vi "Edit Curve.vi"(8 "error in (no error)":errorcluster, 10 "Plot Index":i32, 11 "Data Viewer in":refnum<class "Data Viewer.lvclass">) -> (0 "error out":errorcluster, 1 "Cancel?":bool, 3 "Data Viewer out":refnum<class "Data Viewer.lvclass">)   [LabVIEW 2020, in "Data Viewer.lvlib" / "Data Viewer.lvclass"]
uses:
  Data Viewer.lvclass
  Data Viewer.lvclass/Data Viewer.ctl
panel:
  in  "Tab Control":enum32{"Page 2"}(tab)
  out "名称":string
  in  "Accept":bool
  in  "Data Array":cluster{"Time":timestamp, "Value":dbl}[](array[cluster]) {"Value" format="%.3f"; "Time" format="%<%Y/%m/%d %H:%M:%S%3u>T"}
  in  "Date":timestamp format="%<%Y/%m/%d %H:%M:%S%3u>T"
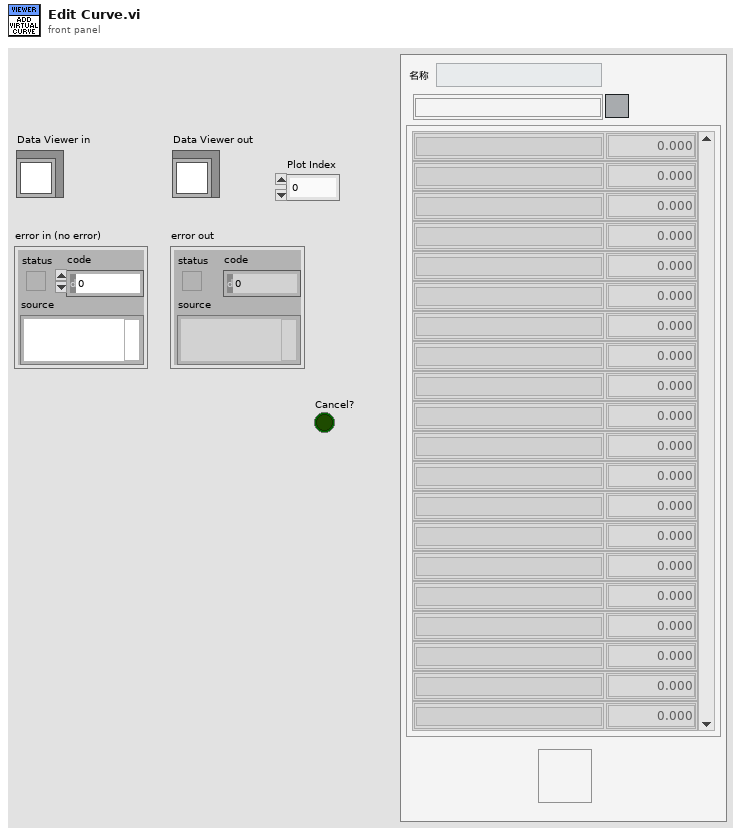
[diagram p1: front panel]
types:
  T1 = enum32{"Invalid", "Standard", "Closed", "Hidden", "Minimized", "Maximized"}
  T2 = typedef "Data Viewer.lvlib/Data Viewer.lvclass/Plot Property--cluster.ctl" = cluster{"Name":string, "Visible":bool, "Color":u32, "Scale Index":i32, "Show Peak Line":bool}
  T3 = typedef "Data Viewer.lvlib/Data Serie--cluster.ctl" = cluster{"Name":string, "Unit":string, "Sample Rate[Hz]":dbl, "Delta t[S]":dbl, "t0":timestamp, "Length":i32, "Time":timestamp[], "Value":dbl[]}
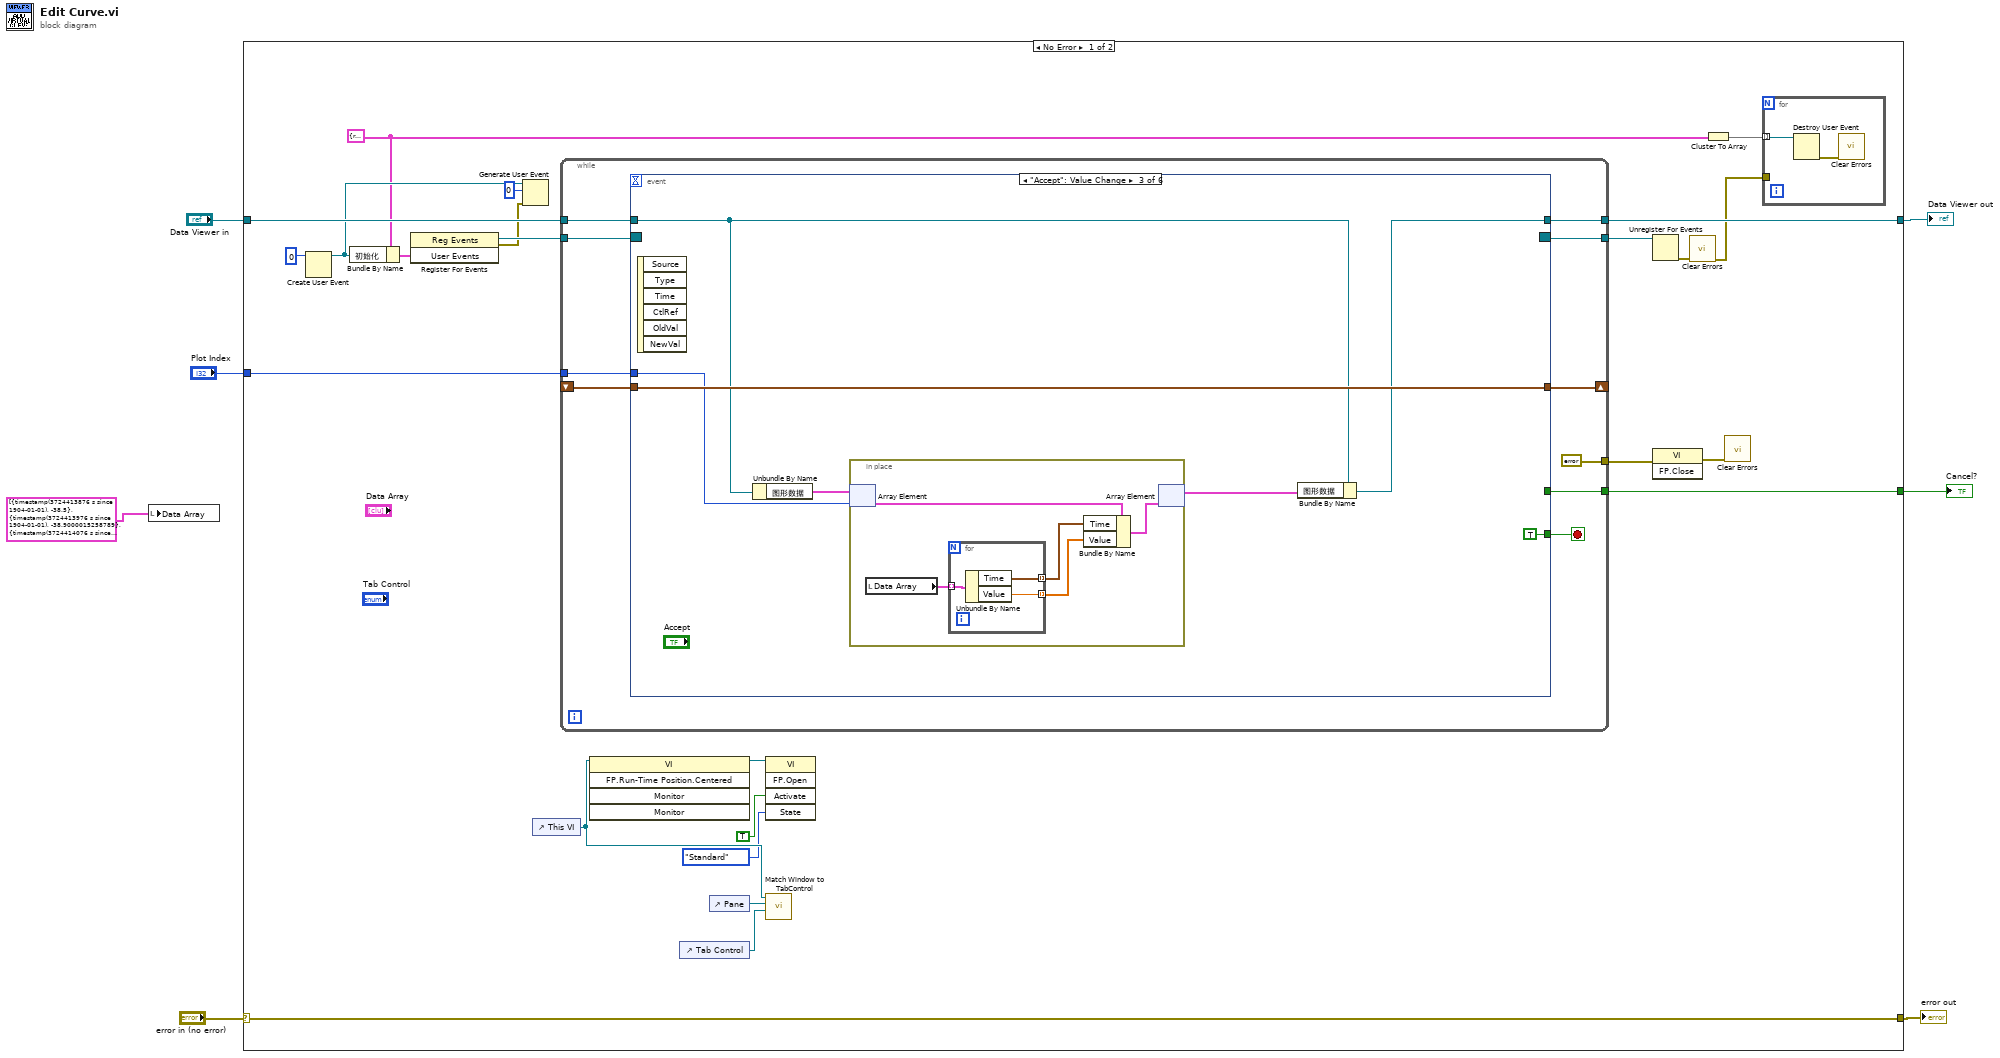
[diagram p0: block diagram]
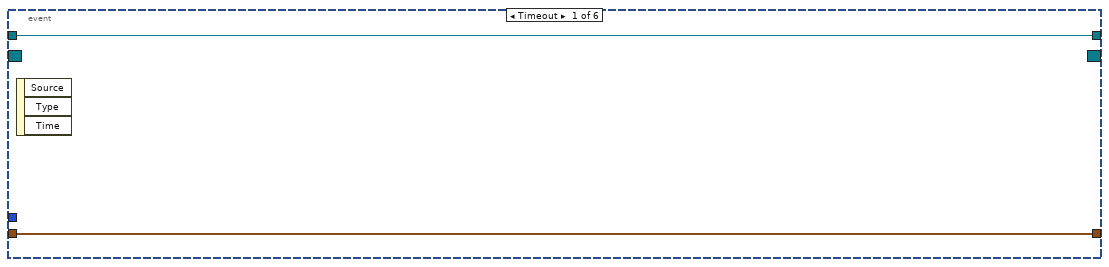
[diagram p2: hidden frame]
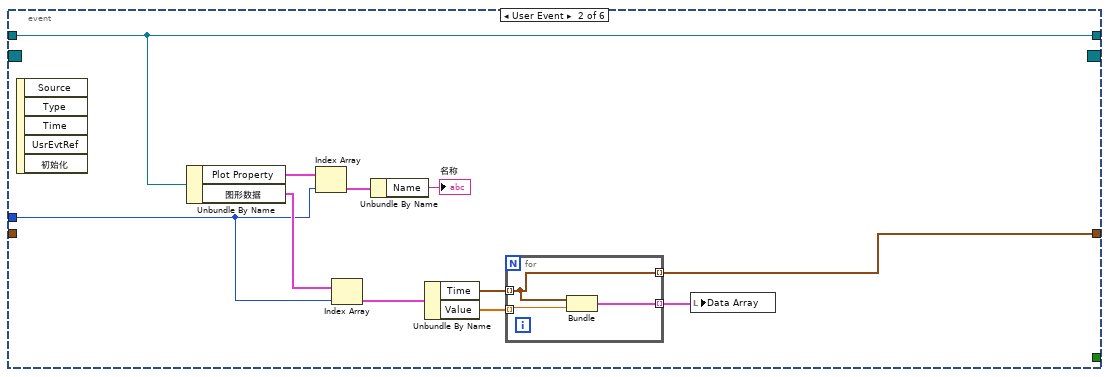
[diagram p3: hidden frame]
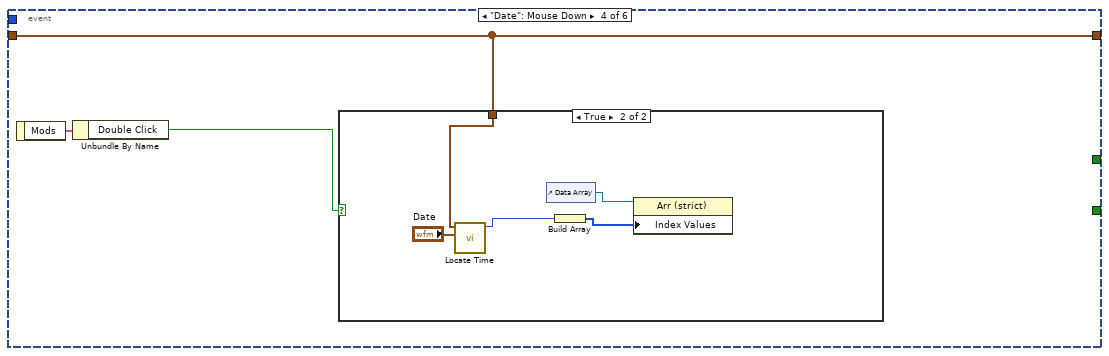
[diagram p4: hidden frame]
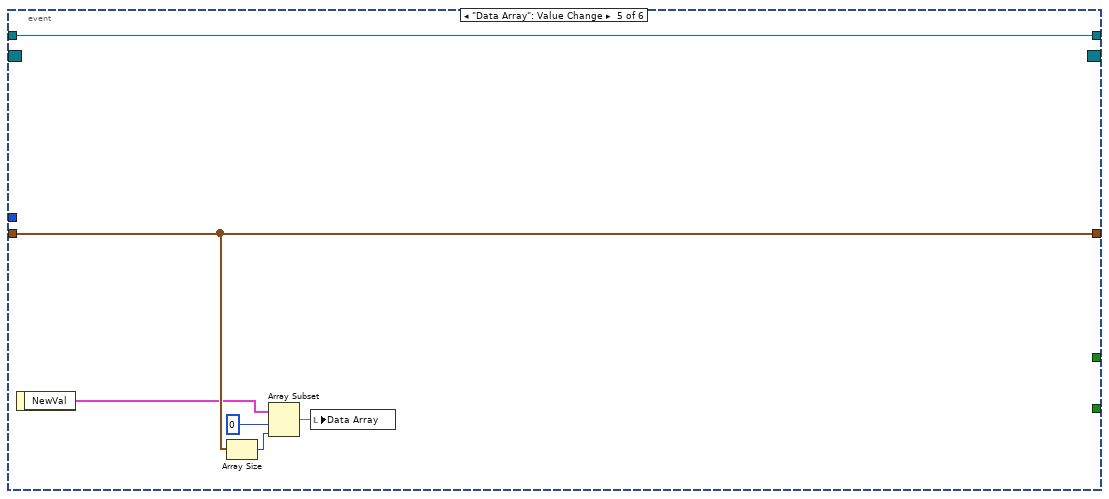
[diagram p6: hidden frame]
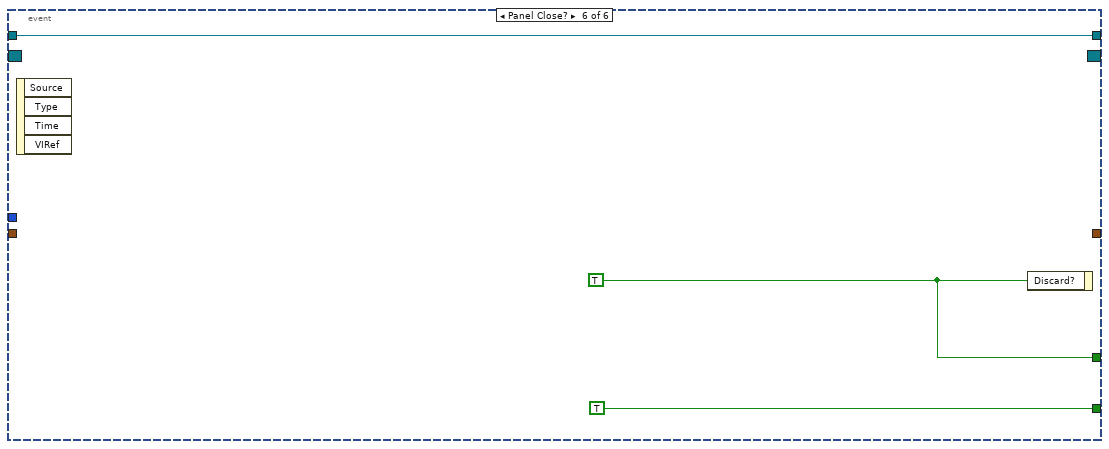
[diagram p7: hidden frame]
diagram:
  n1 = local write "Data Array"(cluster{"数值":timestamp, "数值 2":dbl}[] [{"数值"=timestamp(3724413876.000003 s since 1904-01-01), "数值 2"=-38.5}, {"数值"=timestamp(3724413976.000003 s since 1904-01-01), "数值 2"=-38.9000015258789}, {"数值"=timestamp(3724414076.000003 s since 1904-01-01), "数值 2"=-40.7000007629395}, {"数值"=timestamp(3724414176.000003 s since 1904-01-01), "数值 2"=-41.2000007629395}, {"数值"=timestamp(3724414276.000003 s since 1904-01-01), "数值 2"=-40.5999984741211}, {"数值"=timestamp(3724414376.000003 s since 1904-01-01), "数值 2"=-38.7000007629395}, {"数值"=timestamp(3724414476.000003 s since 1904-01-01), "数值 2"=-38.7000007629395}, {"数值"=timestamp(3724414576.000003 s since 1904-01-01), "数值 2"=-40.4000015258789}, {"数值"=timestamp(3724414676.000003 s since 1904-01-01), "数值 2"=-41.0999984741211}, {"数值"=timestamp(3724414776.000003 s since 1904-01-01), "数值 2"=-40.7999992370605}, {"数值"=timestamp(3724414876.000003 s since 1904-01-01), "数值 2"=-39.5999984741211}, {"数值"=timestamp(3724414976.000003 s since 1904-01-01), "数值 2"=59.5}, {"数值"=timestamp(3724415076.000003 s since 1904-01-01), "数值 2"=86.3000030517578}, {"数值"=timestamp(3724415176.000003 s since 1904-01-01), "数值 2"=85.1999969482422}, {"数值"=timestamp(3724415276.000003 s since 1904-01-01), "数值 2"=85.0999984741211}, {"数值"=timestamp(3724415376.000003 s since 1904-01-01), "数值 2"=85.0}, {"数值"=timestamp(3724415476.000003 s since 1904-01-01), "数值 2"=85.0}, {"数值"=timestamp(3724415576.000003 s since 1904-01-01), "数值 2"=85.0}, {"数值"=timestamp(3724415676.000003 s since 1904-01-01), "数值 2"=85.0}, {"数值"=timestamp(3724415776.000003 s since 1904-01-01), "数值 2"=85.0}, {"数值"=timestamp(3724415876.000003 s since 1904-01-01), "数值 2"=85.0}, {"数值"=timestamp(3724415976.000003 s since 1904-01-01), "数值 2"=85.0}, {"数值"=timestamp(3724416076.000003 s since 1904-01-01), "数值 2"=85.0}, {"数值"=timestamp(3724416176.000003 s since 1904-01-01), "数值 2"=85.0999984741211}, {"数值"=timestamp(3724416276.000003 s since 1904-01-01), "数值 2"=84.9000015258789}, {"数值"=timestamp(3724416376.000003 s since 1904-01-01), "数值 2"=84.9000015258789}, {"数值"=timestamp(3724416476.000003 s since 1904-01-01), "数值 2"=84.9000015258789}, {"数值"=timestamp(3724416576.000003 s since 1904-01-01), "数值 2"=85.0}, {"数值"=timestamp(3724416676.000003 s since 1904-01-01), "数值 2"=85.0}, {"数值"=timestamp(3724416776.000003 s since 1904-01-01), "数值 2"=-2.0}, {"数值"=timestamp(3724416876.000003 s since 1904-01-01), "数值 2"=-42.5}, {"数值"=timestamp(3724416976.000003 s since 1904-01-01), "数值 2"=-40.7999992370605}, {"数值"=timestamp(3724417076.000003 s since 1904-01-01), "数值 2"=-40.2999992370605}, {"数值"=timestamp(3724417176.000003 s since 1904-01-01), "数值 2"=-38.0999984741211}, {"数值"=timestamp(3724417276.000003 s since 1904-01-01), "数值 2"=-38.2000007629395}, {"数值"=timestamp(3724417376.000003 s since 1904-01-01), "数值 2"=-39.0999984741211}, {"数值"=timestamp(3724417476.000003 s since 1904-01-01), "数值 2"=-40.4000015258789}, {"数值"=timestamp(3724417576.000003 s since 1904-01-01), "数值 2"=-41.0}, {"数值"=timestamp(3724417676.000003 s since 1904-01-01), "数值 2"=-41.0}, {"数值"=timestamp(3724417776.000003 s since 1904-01-01), "数值 2"=-39.7000007629395}, {"数值"=timestamp(3724417876.000003 s since 1904-01-01), "数值 2"=-38.5999984741211}, {"数值"=timestamp(3724417976.000003 s since 1904-01-01), "数值 2"=-39.2999992370605}, {"数值"=timestamp(3724418076.000003 s since 1904-01-01), "数值 2"=-40.9000015258789}, {"数值"=timestamp(3724418176.000003 s since 1904-01-01), "数值 2"=-41.2000007629395}, {"数值"=timestamp(3724418276.000003 s since 1904-01-01), "数值 2"=-40.5999984741211}, {"数值"=timestamp(3724418376.000003 s since 1904-01-01), "数值 2"=-38.7999992370605}, {"数值"=timestamp(3724418476.000003 s since 1904-01-01), "数值 2"=-38.5999984741211}, {"数值"=timestamp(3724418576.000003 s since 1904-01-01), "数值 2"=-40.0999984741211}, {"数值"=timestamp(3724418676.000003 s since 1904-01-01), "数值 2"=-41.0999984741211}, {"数值"=timestamp(3724418776.000003 s since 1904-01-01), "数值 2"=-40.9000015258789}, {"数值"=timestamp(3724418876.000003 s since 1904-01-01), "数值 2"=-39.9000015258789}, {"数值"=timestamp(3724418976.000003 s since 1904-01-01), "数值 2"=-38.5999984741211}, {"数值"=timestamp(3724419076.000003 s since 1904-01-01), "数值 2"=-39.5999984741211}, {"数值"=timestamp(3724419176.000003 s since 1904-01-01), "数值 2"=-40.7000007629395}, {"数值"=timestamp(3724419276.000003 s since 1904-01-01), "数值 2"=-41.0999984741211}, {"数值"=timestamp(3724419376.000003 s since 1904-01-01), "数值 2"=-40.4000015258789}, {"数值"=timestamp(3724419476.000003 s since 1904-01-01), "数值 2"=-37.0}, {"数值"=timestamp(3724419576.000003 s since 1904-01-01), "数值 2"=86.4000015258789}, {"数值"=timestamp(3724419676.000003 s since 1904-01-01), "数值 2"=85.0}, {"数值"=timestamp(3724419776.000003 s since 1904-01-01), "数值 2"=85.0999984741211}, {"数值"=timestamp(3724419876.000003 s since 1904-01-01), "数值 2"=85.0}, {"数值"=timestamp(3724419976.000003 s since 1904-01-01), "数值 2"=84.9000015258789}, {"数值"=timestamp(3724420076.000003 s since 1904-01-01), "数值 2"=84.9000015258789}, {"数值"=timestamp(3724420176.000003 s since 1904-01-01), "数值 2"=85.0}, {"数值"=timestamp(3724420276.000003 s since 1904-01-01), "数值 2"=85.0}, {"数值"=timestamp(3724420376.000003 s since 1904-01-01), "数值 2"=85.0999984741211}, {"数值"=timestamp(3724420476.000003 s since 1904-01-01), "数值 2"=84.9000015258789}, {"数值"=timestamp(3724420576.000003 s since 1904-01-01), "数值 2"=84.9000015258789}, {"数值"=timestamp(3724420676.000003 s since 1904-01-01), "数值 2"=85.0}, {"数值"=timestamp(3724420776.000003 s since 1904-01-01), "数值 2"=85.0}, {"数值"=timestamp(3724420876.000003 s since 1904-01-01), "数值 2"=85.0}, {"数值"=timestamp(3724420976.000003 s since 1904-01-01), "数值 2"=84.9000015258789}, {"数值"=timestamp(3724421076.000003 s since 1904-01-01), "数值 2"=85.0999984741211}, {"数值"=timestamp(3724421176.000003 s since 1904-01-01), "数值 2"=85.0}, {"数值"=timestamp(3724421276.000003 s since 1904-01-01), "数值 2"=76.1999969482422}, {"数值"=timestamp(3724421376.000003 s since 1904-01-01), "数值 2"=-42.0999984741211}, {"数值"=timestamp(3724421476.000003 s since 1904-01-01), "数值 2"=-40.7999992370605}, {"数值"=timestamp(3724421576.000003 s since 1904-01-01), "数值 2"=-40.2999992370605}, {"数值"=timestamp(3724421676.000003 s since 1904-01-01), "数值 2"=-38.0}, {"数值"=timestamp(3724421776.000003 s since 1904-01-01), "数值 2"=-38.2999992370605}, {"数值"=timestamp(3724421876.000003 s since 1904-01-01), "数值 2"=-39.0999984741211}, {"数值"=timestamp(3724421976.000003 s since 1904-01-01), "数值 2"=-40.7000007629395}, {"数值"=timestamp(3724422076.000003 s since 1904-01-01), "数值 2"=-41.2000007629395}, {"数值"=timestamp(3724422176.000003 s since 1904-01-01), "数值 2"=-40.9000015258789}, {"数值"=timestamp(3724422276.000003 s since 1904-01-01), "数值 2"=-39.2999992370605}, {"数值"=timestamp(3724422376.000003 s since 1904-01-01), "数值 2"=-38.7000007629395}, {"数值"=timestamp(3724422476.000003 s since 1904-01-01), "数值 2"=-39.9000015258789}, {"数值"=timestamp(3724422576.000003 s since 1904-01-01), "数值 2"=-41.0}, {"数值"=timestamp(3724422676.000003 s since 1904-01-01), "数值 2"=-41.0}, {"数值"=timestamp(3724422776.000003 s since 1904-01-01), "数值 2"=-40.2000007629395}, {"数值"=timestamp(3724422876.000003 s since 1904-01-01), "数值 2"=-38.5999984741211}, {"数值"=timestamp(3724422976.000003 s since 1904-01-01), "数值 2"=-39.0}, {"数值"=timestamp(3724423076.000003 s since 1904-01-01), "数值 2"=-40.5}, {"数值"=timestamp(3724423176.000003 s since 1904-01-01), "数值 2"=-41.2000007629395}, {"数值"=timestamp(3724423276.000003 s since 1904-01-01), "数值 2"=-40.7999992370605}, {"数值"=timestamp(3724423376.000003 s since 1904-01-01), "数值 2"=-39.5999984741211}, {"数值"=timestamp(3724423476.000003 s since 1904-01-01), "数值 2"=-38.5999984741211}, {"数值"=timestamp(3724423576.000003 s since 1904-01-01), "数值 2"=-39.7999992370605}, {"数值"=timestamp(3724423676.000003 s since 1904-01-01), "数值 2"=-40.7999992370605}, {"数值"=timestamp(3724423776.000003 s since 1904-01-01), "数值 2"=-41.0}, {"数值"=timestamp(3724423876.000003 s since 1904-01-01), "数值 2"=-40.2000007629395}, {"数值"=timestamp(3724423976.000003 s since 1904-01-01), "数值 2"=-6.90000009536743}, {"数值"=timestamp(3724424076.000003 s since 1904-01-01), "数值 2"=86.0}, {"数值"=timestamp(3724424176.000003 s since 1904-01-01), "数值 2"=85.0999984741211}, {"数值"=timestamp(3724424276.000003 s since 1904-01-01), "数值 2"=85.0}, {"数值"=timestamp(3724424376.000003 s since 1904-01-01), "数值 2"=85.0}, {"数值"=timestamp(3724424476.000003 s since 1904-01-01), "数值 2"=85.0}, {"数值"=timestamp(3724424576.000003 s since 1904-01-01), "数值 2"=85.0}, {"数值"=timestamp(3724424676.000003 s since 1904-01-01), "数值 2"=85.0}, {"数值"=timestamp(3724424776.000003 s since 1904-01-01), "数值 2"=85.0}, {"数值"=timestamp(3724424876.000003 s since 1904-01-01), "数值 2"=85.0}, {"数值"=timestamp(3724424976.000003 s since 1904-01-01), "数值 2"=85.0}, {"数值"=timestamp(3724425076.000003 s since 1904-01-01), "数值 2"=84.9000015258789}, {"数值"=timestamp(3724425176.000003 s since 1904-01-01), "数值 2"=84.9000015258789}, {"数值"=timestamp(3724425276.000003 s since 1904-01-01), "数值 2"=85.0999984741211}, {"数值"=timestamp(3724425376.000003 s since 1904-01-01), "数值 2"=84.9000015258789}, {"数值"=timestamp(3724425476.000003 s since 1904-01-01), "数值 2"=85.0}, {"数值"=timestamp(3724425576.000003 s since 1904-01-01), "数值 2"=85.0999984741211}, {"数值"=timestamp(3724425676.000003 s since 1904-01-01), "数值 2"=84.9000015258789}, {"数值"=timestamp(3724425776.000003 s since 1904-01-01), "数值 2"=47.9000015258789}, {"数值"=timestamp(3724425876.000003 s since 1904-01-01), "数值 2"=-43.7000007629395}, {"数值"=timestamp(3724425976.000003 s since 1904-01-01), "数值 2"=-40.5999984741211}, {"数值"=timestamp(3724426076.000003 s since 1904-01-01), "数值 2"=-40.2999992370605}, {"数值"=timestamp(3724426176.000003 s since 1904-01-01), "数值 2"=-38.5}, {"数值"=timestamp(3724426276.000003 s since 1904-01-01), "数值 2"=-38.2999992370605}, {"数值"=timestamp(3724426376.000003 s since 1904-01-01), "数值 2"=-39.0}, {"数值"=timestamp(3724426476.000003 s since 1904-01-01), "数值 2"=-40.4000015258789}, {"数值"=timestamp(3724426576.000003 s since 1904-01-01), "数值 2"=-41.0999984741211}, {"数值"=timestamp(3724426676.000003 s since 1904-01-01), "数值 2"=-40.7999992370605}, {"数值"=timestamp(3724426776.000003 s since 1904-01-01), "数值 2"=-39.5999984741211}, {"数值"=timestamp(3724426876.000003 s since 1904-01-01), "数值 2"=-38.7000007629395}, {"数值"=timestamp(3724426976.000003 s since 1904-01-01), "数值 2"=-40.0999984741211}, {"数值"=timestamp(3724427076.000003 s since 1904-01-01), "数值 2"=-40.7000007629395}, {"数值"=timestamp(3724427176.000003 s since 1904-01-01), "数值 2"=-40.7999992370605}, {"数值"=timestamp(3724427276.000003 s since 1904-01-01), "数值 2"=-39.9000015258789}, {"数值"=timestamp(3724427376.000003 s since 1904-01-01), "数值 2"=-38.7000007629395}, {"数值"=timestamp(3724427476.000003 s since 1904-01-01), "数值 2"=-39.7000007629395}, {"数值"=timestamp(3724427576.000003 s since 1904-01-01), "数值 2"=-40.7999992370605}, {"数值"=timestamp(3724427676.000003 s since 1904-01-01), "数值 2"=-41.0999984741211}, {"数值"=timestamp(3724427776.000003 s since 1904-01-01), "数值 2"=-40.2999992370605}, {"数值"=timestamp(3724427876.000003 s since 1904-01-01), "数值 2"=-39.0}, {"数值"=timestamp(3724427976.000003 s since 1904-01-01), "数值 2"=-38.7000007629395}, {"数值"=timestamp(3724428076.000003 s since 1904-01-01), "数值 2"=-40.4000015258789}, {"数值"=timestamp(3724428176.000003 s since 1904-01-01), "数值 2"=-41.0999984741211}, {"数值"=timestamp(3724428276.000003 s since 1904-01-01), "数值 2"=-40.7999992370605}, {"数值"=timestamp(3724428376.000003 s since 1904-01-01), "数值 2"=-39.5}, {"数值"=timestamp(3724428476.000003 s since 1904-01-01), "数值 2"=25.3999996185303}, {"数值"=timestamp(3724428576.000003 s since 1904-01-01), "数值 2"=86.4000015258789}, {"数值"=timestamp(3724428676.000003 s since 1904-01-01), "数值 2"=85.0999984741211}, {"数值"=timestamp(3724428776.000003 s since 1904-01-01), "数值 2"=85.0}, {"数值"=timestamp(3724428876.000003 s since 1904-01-01), "数值 2"=84.9000015258789}, {"数值"=timestamp(3724428976.000003 s since 1904-01-01), "数值 2"=85.0}, {"数值"=timestamp(3724429076.000003 s since 1904-01-01), "数值 2"=85.0}, {"数值"=timestamp(3724429176.000003 s since 1904-01-01), "数值 2"=85.0}, {"数值"=timestamp(3724429276.000003 s since 1904-01-01), "数值 2"=85.0}, {"数值"=timestamp(3724429376.000003 s since 1904-01-01), "数值 2"=85.0}, {"数值"=timestamp(3724429476.000003 s since 1904-01-01), "数值 2"=85.0}, {"数值"=timestamp(3724429576.000003 s since 1904-01-01), "数值 2"=85.0}, {"数值"=timestamp(3724429676.000003 s since 1904-01-01), "数值 2"=85.0}, {"数值"=timestamp(3724429776.000003 s since 1904-01-01), "数值 2"=85.0999984741211}, {"数值"=timestamp(3724429876.000003 s since 1904-01-01), "数值 2"=84.9000015258789}, {"数值"=timestamp(3724429976.000003 s since 1904-01-01), "数值 2"=85.0}, {"数值"=timestamp(3724430076.000003 s since 1904-01-01), "数值 2"=85.0}, {"数值"=timestamp(3724430176.000003 s since 1904-01-01), "数值 2"=85.0}, {"数值"=timestamp(3724430276.000003 s since 1904-01-01), "数值 2"=18.2000007629395}, {"数值"=timestamp(3724430376.000003 s since 1904-01-01), "数值 2"=-42.7999992370605}, {"数值"=timestamp(3724430476.000003 s since 1904-01-01), "数值 2"=-40.5999984741211}, {"数值"=timestamp(3724430576.000003 s since 1904-01-01), "数值 2"=-40.2000007629395}, {"数值"=timestamp(3724430676.000003 s since 1904-01-01), "数值 2"=-38.2000007629395}, {"数值"=timestamp(3724430776.000003 s since 1904-01-01), "数值 2"=-38.4000015258789}, {"数值"=timestamp(3724430876.000003 s since 1904-01-01), "数值 2"=-39.0999984741211}, {"数值"=timestamp(3724430976.000003 s since 1904-01-01), "数值 2"=-40.5}, {"数值"=timestamp(3724431076.000003 s since 1904-01-01), "数值 2"=-41.0}, {"数值"=timestamp(3724431176.000003 s since 1904-01-01), "数值 2"=-40.5999984741211}, {"数值"=timestamp(3724431276.000003 s since 1904-01-01), "数值 2"=-39.5}, {"数值"=timestamp(3724431376.000003 s since 1904-01-01), "数值 2"=-38.7999992370605}, {"数值"=timestamp(3724431476.000003 s since 1904-01-01), "数值 2"=-40.0}, {"数值"=timestamp(3724431576.000003 s since 1904-01-01), "数值 2"=-40.9000015258789}, {"数值"=timestamp(3724431676.000003 s since 1904-01-01), "数值 2"=-41.0999984741211}, {"数值"=timestamp(3724431776.000003 s since 1904-01-01), "数值 2"=-40.0}, {"数值"=timestamp(3724431876.000003 s since 1904-01-01), "数值 2"=-38.7000007629395}, {"数值"=timestamp(3724431976.000003 s since 1904-01-01), "数值 2"=-38.9000015258789}, {"数值"=timestamp(3724432076.000003 s since 1904-01-01), "数值 2"=-40.5999984741211}, {"数值"=timestamp(3724432176.000003 s since 1904-01-01), "数值 2"=-41.0999984741211}, {"数值"=timestamp(3724432276.000003 s since 1904-01-01), "数值 2"=-40.9000015258789}, {"数值"=timestamp(3724432376.000003 s since 1904-01-01), "数值 2"=-39.5999984741211}, {"数值"=timestamp(3724432476.000003 s since 1904-01-01), "数值 2"=-38.5999984741211}, {"数值"=timestamp(3724432576.000003 s since 1904-01-01), "数值 2"=-39.2999992370605}, {"数值"=timestamp(3724432676.000003 s since 1904-01-01), "数值 2"=-40.9000015258789}, {"数值"=timestamp(3724432776.000003 s since 1904-01-01), "数值 2"=-41.0}, {"数值"=timestamp(3724432876.000003 s since 1904-01-01), "数值 2"=-40.5}, {"数值"=timestamp(3724432976.000003 s since 1904-01-01), "数值 2"=54.9000015258789}, {"数值"=timestamp(3724433076.000003 s since 1904-01-01), "数值 2"=86.5}, {"数值"=timestamp(3724433176.000003 s since 1904-01-01), "数值 2"=85.1999969482422}, {"数值"=timestamp(3724433276.000003 s since 1904-01-01), "数值 2"=85.0999984741211}, {"数值"=timestamp(3724433376.000003 s since 1904-01-01), "数值 2"=85.0}, {"数值"=timestamp(3724433476.000003 s since 1904-01-01), "数值 2"=85.0}, {"数值"=timestamp(3724433576.000003 s since 1904-01-01), "数值 2"=85.0}, {"数值"=timestamp(3724433676.000003 s since 1904-01-01), "数值 2"=85.0}, {"数值"=timestamp(3724433776.000003 s since 1904-01-01), "数值 2"=85.0}, {"数值"=timestamp(3724433876.000003 s since 1904-01-01), "数值 2"=84.9000015258789}, {"数值"=timestamp(3724433976.000003 s since 1904-01-01), "数值 2"=85.0}, {"数值"=timestamp(3724434076.000003 s since 1904-01-01), "数值 2"=85.0999984741211}, {"数值"=timestamp(3724434176.000003 s since 1904-01-01), "数值 2"=85.0}, {"数值"=timestamp(3724434276.000003 s since 1904-01-01), "数值 2"=85.0999984741211}, {"数值"=timestamp(3724434376.000003 s since 1904-01-01), "数值 2"=85.0999984741211}, {"数值"=timestamp(3724434476.000003 s since 1904-01-01), "数值 2"=85.0}, {"数值"=timestamp(3724434576.000003 s since 1904-01-01), "数值 2"=85.0999984741211}, {"数值"=timestamp(3724434676.000003 s since 1904-01-01), "数值 2"=85.0}, {"数值"=timestamp(3724434776.000003 s since 1904-01-01), "数值 2"=3.20000004768372}, {"数值"=timestamp(3724434876.000003 s since 1904-01-01), "数值 2"=-42.7999992370605}, {"数值"=timestamp(3724434976.000003 s since 1904-01-01), "数值 2"=-41.0}, {"数值"=timestamp(3724435076.000003 s since 1904-01-01), "数值 2"=-40.2999992370605}, {"数值"=timestamp(3724435176.000003 s since 1904-01-01), "数值 2"=-38.0999984741211}, {"数值"=timestamp(3724435276.000003 s since 1904-01-01), "数值 2"=-38.2000007629395}, {"数值"=timestamp(3724435376.000003 s since 1904-01-01), "数值 2"=-39.2000007629395}, {"数值"=timestamp(3724435476.000003 s since 1904-01-01), "数值 2"=-40.5}, {"数值"=timestamp(3724435576.000003 s since 1904-01-01), "数值 2"=-41.0999984741211}, {"数值"=timestamp(3724435676.000003 s since 1904-01-01), "数值 2"=-40.7000007629395}, {"数值"=timestamp(3724435776.000003 s since 1904-01-01), "数值 2"=-39.5999984741211}, {"数值"=timestamp(3724435876.000003 s since 1904-01-01), "数值 2"=-38.5999984741211}, {"数值"=timestamp(3724435976.000003 s since 1904-01-01), "数值 2"=-40.0}, {"数值"=timestamp(3724436076.000003 s since 1904-01-01), "数值 2"=-40.9000015258789}, {"数值"=timestamp(3724436176.000003 s since 1904-01-01), "数值 2"=-41.0999984741211}, {"数值"=timestamp(3724436276.000003 s since 1904-01-01), "数值 2"=-40.0}, {"数值"=timestamp(3724436376.000003 s since 1904-01-01), "数值 2"=-38.7000007629395}, {"数值"=timestamp(3724436476.000003 s since 1904-01-01), "数值 2"=-38.9000015258789}, {"数值"=timestamp(3724436576.000003 s since 1904-01-01), "数值 2"=-40.5999984741211}, {"数值"=timestamp(3724436676.000003 s since 1904-01-01), "数值 2"=-41.2000007629395}, {"数值"=timestamp(3724436776.000003 s since 1904-01-01), "数值 2"=-40.9000015258789}, {"数值"=timestamp(3724436876.000003 s since 1904-01-01), "数值 2"=-39.5}, {"数值"=timestamp(3724436976.000003 s since 1904-01-01), "数值 2"=-38.5999984741211}, {"数值"=timestamp(3724437076.000003 s since 1904-01-01), "数值 2"=-39.5}, {"数值"=timestamp(3724437176.000003 s since 1904-01-01), "数值 2"=-40.9000015258789}, {"数值"=timestamp(3724437276.000003 s since 1904-01-01), "数值 2"=-41.0}, {"数值"=timestamp(3724437376.000003 s since 1904-01-01), "数值 2"=-40.2999992370605}, {"数值"=timestamp(3724437476.000003 s since 1904-01-01), "数值 2"=71.5999984741211}, {"数值"=timestamp(3724437576.000003 s since 1904-01-01), "数值 2"=86.4000015258789}, {"数值"=timestamp(3724437676.000003 s since 1904-01-01), "数值 2"=85.0}, {"数值"=timestamp(3724437776.000003 s since 1904-01-01), "数值 2"=85.0999984741211}, {"数值"=timestamp(3724437876.000003 s since 1904-01-01), "数值 2"=85.0}, {"数值"=timestamp(3724437976.000003 s since 1904-01-01), "数值 2"=85.0}, {"数值"=timestamp(3724438076.000003 s since 1904-01-01), "数值 2"=85.0}, {"数值"=timestamp(3724438176.000003 s since 1904-01-01), "数值 2"=85.0}, {"数值"=timestamp(3724438276.000003 s since 1904-01-01), "数值 2"=85.0}, {"数值"=timestamp(3724438376.000003 s since 1904-01-01), "数值 2"=85.0}, {"数值"=timestamp(3724438476.000003 s since 1904-01-01), "数值 2"=85.0}, {"数值"=timestamp(3724438576.000003 s since 1904-01-01), "数值 2"=84.9000015258789}, {"数值"=timestamp(3724438676.000003 s since 1904-01-01), "数值 2"=85.0}, {"数值"=timestamp(3724438776.000003 s since 1904-01-01), "数值 2"=85.0999984741211}, {"数值"=timestamp(3724438876.000003 s since 1904-01-01), "数值 2"=85.0}, {"数值"=timestamp(3724438976.000003 s since 1904-01-01), "数值 2"=85.0}, {"数值"=timestamp(3724439076.000003 s since 1904-01-01), "数值 2"=85.0}, {"数值"=timestamp(3724439176.000003 s since 1904-01-01), "数值 2"=85.0999984741211}, {"数值"=timestamp(3724439276.000003 s since 1904-01-01), "数值 2"=79.5}, {"数值"=timestamp(3724439376.000003 s since 1904-01-01), "数值 2"=-42.5999984741211}, {"数值"=timestamp(3724439476.000003 s since 1904-01-01), "数值 2"=-40.9000015258789}, {"数值"=timestamp(3724439576.000003 s since 1904-01-01), "数值 2"=-40.4000015258789}, {"数值"=timestamp(3724439676.000003 s since 1904-01-01), "数值 2"=-38.0999984741211}, {"数值"=timestamp(3724439776.000003 s since 1904-01-01), "数值 2"=-38.2999992370605}, {"数值"=timestamp(3724439876.000003 s since 1904-01-01), "数值 2"=-39.2000007629395}, {"数值"=timestamp(3724439976.000003 s since 1904-01-01), "数值 2"=-40.7999992370605}, {"数值"=timestamp(3724440076.000003 s since 1904-01-01), "数值 2"=-41.0999984741211}, {"数值"=timestamp(3724440176.000003 s since 1904-01-01), "数值 2"=-40.7000007629395}, {"数值"=timestamp(3724440276.000003 s since 1904-01-01), "数值 2"=-38.7999992370605}, {"数值"=timestamp(3724440376.000003 s since 1904-01-01), "数值 2"=-38.9000015258789}, {"数值"=timestamp(3724440476.000003 s since 1904-01-01), "数值 2"=-40.0999984741211}, {"数值"=timestamp(3724440576.000003 s since 1904-01-01), "数值 2"=-41.0}, {"数值"=timestamp(3724440676.000003 s since 1904-01-01), "数值 2"=-40.9000015258789}, {"数值"=timestamp(3724440776.000003 s since 1904-01-01), "数值 2"=-39.9000015258789}, {"数值"=timestamp(3724440876.000003 s since 1904-01-01), "数值 2"=-38.7000007629395}, {"数值"=timestamp(3724440976.000003 s since 1904-01-01), "数值 2"=-39.5}, {"数值"=timestamp(3724441076.000003 s since 1904-01-01), "数值 2"=-40.7999992370605}, {"数值"=timestamp(3724441176.000003 s since 1904-01-01), "数值 2"=-41.0999984741211}, {"数值"=timestamp(3724441276.000003 s since 1904-01-01), "数值 2"=-40.2999992370605}, {"数值"=timestamp(3724441376.000003 s since 1904-01-01), "数值 2"=-38.7999992370605}, {"数值"=timestamp(3724441476.000003 s since 1904-01-01), "数值 2"=-39.0999984741211}, {"数值"=timestamp(3724441576.000003 s since 1904-01-01), "数值 2"=-40.5999984741211}, {"数值"=timestamp(3724441676.000003 s since 1904-01-01), "数值 2"=-41.0}, {"数值"=timestamp(3724441776.000003 s since 1904-01-01), "数值 2"=-40.5}, {"数值"=timestamp(3724441876.000003 s since 1904-01-01), "数值 2"=-39.0}, {"数值"=timestamp(3724441976.000003 s since 1904-01-01), "数值 2"=-23.6000003814697}, {"数值"=timestamp(3724442076.000003 s since 1904-01-01), "数值 2"=86.0999984741211}, {"数值"=timestamp(3724442176.000003 s since 1904-01-01), "数值 2"=85.0}, {"数值"=timestamp(3724442276.000003 s since 1904-01-01), "数值 2"=85.0}, {"数值"=timestamp(3724442376.000003 s since 1904-01-01), "数值 2"=85.0999984741211}, {"数值"=timestamp(3724442476.000003 s since 1904-01-01), "数值 2"=85.0}, {"数值"=timestamp(3724442576.000003 s since 1904-01-01), "数值 2"=85.0}, {"数值"=timestamp(3724442676.000003 s since 1904-01-01), "数值 2"=85.0}, {"数值"=timestamp(3724442776.000003 s since 1904-01-01), "数值 2"=85.0}, {"数值"=timestamp(3724442876.000003 s since 1904-01-01), "数值 2"=85.0}, {"数值"=timestamp(3724442976.000003 s since 1904-01-01), "数值 2"=85.0}, {"数值"=timestamp(3724443076.000003 s since 1904-01-01), "数值 2"=85.0999984741211}, {"数值"=timestamp(3724443176.000003 s since 1904-01-01), "数值 2"=85.0999984741211}, {"数值"=timestamp(3724443276.000003 s since 1904-01-01), "数值 2"=85.0}, {"数值"=timestamp(3724443376.000003 s since 1904-01-01), "数值 2"=85.0999984741211}, {"数值"=timestamp(3724443476.000003 s since 1904-01-01), "数值 2"=85.0}, {"数值"=timestamp(3724443576.000003 s since 1904-01-01), "数值 2"=85.0999984741211}, {"数值"=timestamp(3724443676.000003 s since 1904-01-01), "数值 2"=85.0999984741211}, {"数值"=timestamp(3724443776.000003 s since 1904-01-01), "数值 2"=56.7000007629395}, {"数值"=timestamp(3724443876.000003 s since 1904-01-01), "数值 2"=-42.4000015258789}, {"数值"=timestamp(3724443976.000003 s since 1904-01-01), "数值 2"=-41.2999992370605}, {"数值"=timestamp(3724444076.000003 s since 1904-01-01), "数值 2"=-40.5}, {"数值"=timestamp(3724444176.000003 s since 1904-01-01), "数值 2"=-38.0}, {"数值"=timestamp(3724444276.000003 s since 1904-01-01), "数值 2"=-38.2999992370605}, {"数值"=timestamp(3724444376.000003 s since 1904-01-01), "数值 2"=-39.5}, {"数值"=timestamp(3724444476.000003 s since 1904-01-01), "数值 2"=-40.4000015258789}, {"数值"=timestamp(3724444576.000003 s since 1904-01-01), "数值 2"=-40.7999992370605}, {"数值"=timestamp(3724444676.000003 s since 1904-01-01), "数值 2"=-40.9000015258789}, {"数值"=timestamp(3724444776.000003 s since 1904-01-01), "数值 2"=-39.5999984741211}, {"数值"=timestamp(3724444876.000003 s since 1904-01-01), "数值 2"=-38.5999984741211}, {"数值"=timestamp(3724444976.000003 s since 1904-01-01), "数值 2"=-39.7000007629395}, {"数值"=timestamp(3724445076.000003 s since 1904-01-01), "数值 2"=-40.9000015258789}, {"数值"=timestamp(3724445176.000003 s since 1904-01-01), "数值 2"=-41.0999984741211}, {"数值"=timestamp(3724445276.000003 s since 1904-01-01), "数值 2"=-40.4000015258789}, {"数值"=timestamp(3724445376.000003 s since 1904-01-01), "数值 2"=-38.5999984741211}, {"数值"=timestamp(3724445476.000003 s since 1904-01-01), "数值 2"=-38.9000015258789}, {"数值"=timestamp(3724445576.000003 s since 1904-01-01), "数值 2"=-40.5}, {"数值"=timestamp(3724445676.000003 s since 1904-01-01), "数值 2"=-41.2000007629395}, {"数值"=timestamp(3724445776.000003 s since 1904-01-01), "数值 2"=-40.7999992370605}, {"数值"=timestamp(3724445876.000003 s since 1904-01-01), "数值 2"=-39.5999984741211}, {"数值"=timestamp(3724445976.000003 s since 1904-01-01), "数值 2"=-38.5}, {"数值"=timestamp(3724446076.000003 s since 1904-01-01), "数值 2"=-39.5999984741211}, {"数值"=timestamp(3724446176.000003 s since 1904-01-01), "数值 2"=-40.7999992370605}, {"数值"=timestamp(3724446276.000003 s since 1904-01-01), "数值 2"=-41.0999984741211}, {"数值"=timestamp(3724446376.000003 s since 1904-01-01), "数值 2"=-40.2000007629395}, {"数值"=timestamp(3724446476.000003 s since 1904-01-01), "数值 2"=19.6000003814697}, {"数值"=timestamp(3724446576.000003 s since 1904-01-01), "数值 2"=86.0999984741211}, {"数值"=timestamp(3724446676.000003 s since 1904-01-01), "数值 2"=85.0}, {"数值"=timestamp(3724446776.000003 s since 1904-01-01), "数值 2"=85.0}, {"数值"=timestamp(3724446876.000003 s since 1904-01-01), "数值 2"=85.0}, {"数值"=timestamp(3724446976.000003 s since 1904-01-01), "数值 2"=84.9000015258789}, {"数值"=timestamp(3724447076.000003 s since 1904-01-01), "数值 2"=85.0}, {"数值"=timestamp(3724447176.000003 s since 1904-01-01), "数值 2"=85.0}, {"数值"=timestamp(3724447276.000003 s since 1904-01-01), "数值 2"=85.0}, {"数值"=timestamp(3724447376.000003 s since 1904-01-01), "数值 2"=85.0}, {"数值"=timestamp(3724447476.000003 s since 1904-01-01), "数值 2"=85.0}, {"数值"=timestamp(3724447576.000003 s since 1904-01-01), "数值 2"=85.0}, {"数值"=timestamp(3724447676.000003 s since 1904-01-01), "数值 2"=85.0}, {"数值"=timestamp(3724447776.000003 s since 1904-01-01), "数值 2"=85.0}, {"数值"=timestamp(3724447876.000003 s since 1904-01-01), "数值 2"=85.0}, {"数值"=timestamp(3724447976.000003 s since 1904-01-01), "数值 2"=85.0}, {"数值"=timestamp(3724448076.000003 s since 1904-01-01), "数值 2"=85.0}, {"数值"=timestamp(3724448176.000003 s since 1904-01-01), "数值 2"=85.0}, {"数值"=timestamp(3724448276.000003 s since 1904-01-01), "数值 2"=25.1000003814697}, {"数值"=timestamp(3724448376.000003 s since 1904-01-01), "数值 2"=-43.5}, {"数值"=timestamp(3724448476.000003 s since 1904-01-01), "数值 2"=-40.9000015258789}, {"数值"=timestamp(3724448576.000003 s since 1904-01-01), "数值 2"=-40.2999992370605}, {"数值"=timestamp(3724448676.000003 s since 1904-01-01), "数值 2"=-38.0999984741211}, {"数值"=timestamp(3724448776.000003 s since 1904-01-01), "数值 2"=-38.2999992370605}, {"数值"=timestamp(3724448876.000003 s since 1904-01-01), "数值 2"=-39.0999984741211}, {"数值"=timestamp(3724448976.000003 s since 1904-01-01), "数值 2"=-40.4000015258789}, {"数值"=timestamp(3724449076.000003 s since 1904-01-01), "数值 2"=-41.2000007629395}, {"数值"=timestamp(3724449176.000003 s since 1904-01-01), "数值 2"=-40.7999992370605}, {"数值"=timestamp(3724449276.000003 s since 1904-01-01), "数值 2"=-39.5}, {"数值"=timestamp(3724449376.000003 s since 1904-01-01), "数值 2"=-38.7000007629395}, {"数值"=timestamp(3724449476.000003 s since 1904-01-01), "数值 2"=-40.0999984741211}, {"数值"=timestamp(3724449576.000003 s since 1904-01-01), "数值 2"=-40.9000015258789}, {"数值"=timestamp(3724449676.000003 s since 1904-01-01), "数值 2"=-40.7999992370605}, {"数值"=timestamp(3724449776.000003 s since 1904-01-01), "数值 2"=-39.7999992370605}, {"数值"=timestamp(3724449876.000003 s since 1904-01-01), "数值 2"=-38.5999984741211}, {"数值"=timestamp(3724449976.000003 s since 1904-01-01), "数值 2"=-39.5999984741211}, {"数值"=timestamp(3724450076.000003 s since 1904-01-01), "数值 2"=-40.7999992370605}, {"数值"=timestamp(3724450176.000003 s since 1904-01-01), "数值 2"=-41.2000007629395}, {"数值"=timestamp(3724450276.000003 s since 1904-01-01), "数值 2"=-40.2999992370605}, {"数值"=timestamp(3724450376.000003 s since 1904-01-01), "数值 2"=-38.9000015258789}, {"数值"=timestamp(3724450476.000003 s since 1904-01-01), "数值 2"=-38.7000007629395}, {"数值"=timestamp(3724450576.000003 s since 1904-01-01), "数值 2"=-40.4000015258789}, {"数值"=timestamp(3724450676.000003 s since 1904-01-01), "数值 2"=-41.2999992370605}, {"数值"=timestamp(3724450776.000003 s since 1904-01-01), "数值 2"=-41.0}, {"数值"=timestamp(3724450876.000003 s since 1904-01-01), "数值 2"=-39.5}, {"数值"=timestamp(3724450976.000003 s since 1904-01-01), "数值 2"=46.5999984741211}, {"数值"=timestamp(3724451076.000003 s since 1904-01-01), "数值 2"=86.1999969482422}, {"数值"=timestamp(3724451176.000003 s since 1904-01-01), "数值 2"=85.1999969482422}, {"数值"=timestamp(3724451276.000003 s since 1904-01-01), "数值 2"=85.0999984741211}, {"数值"=timestamp(3724451376.000003 s since 1904-01-01), "数值 2"=85.0999984741211}, {"数值"=timestamp(3724451476.000003 s since 1904-01-01), "数值 2"=85.0}, {"数值"=timestamp(3724451576.000003 s since 1904-01-01), "数值 2"=84.9000015258789}, {"数值"=timestamp(3724451676.000003 s since 1904-01-01), "数值 2"=85.0}, {"数值"=timestamp(3724451776.000003 s since 1904-01-01), "数值 2"=85.0}, {"数值"=timestamp(3724451876.000003 s since 1904-01-01), "数值 2"=85.0999984741211}, {"数值"=timestamp(3724451976.000003 s since 1904-01-01), "数值 2"=85.0}, {"数值"=timestamp(3724452076.000003 s since 1904-01-01), "数值 2"=84.9000015258789}, {"数值"=timestamp(3724452176.000003 s since 1904-01-01), "数值 2"=85.0}, {"数值"=timestamp(3724452276.000003 s since 1904-01-01), "数值 2"=84.9000015258789}, {"数值"=timestamp(3724452376.000003 s since 1904-01-01), "数值 2"=85.0}, {"数值"=timestamp(3724452476.000003 s since 1904-01-01), "数值 2"=85.0999984741211}, {"数值"=timestamp(3724452576.000003 s since 1904-01-01), "数值 2"=85.0}, {"数值"=timestamp(3724452676.000003 s since 1904-01-01), "数值 2"=85.0}, {"数值"=timestamp(3724452776.000003 s since 1904-01-01), "数值 2"=3.90000009536743}, {"数值"=timestamp(3724452876.000003 s since 1904-01-01), "数值 2"=-43.0}, {"数值"=timestamp(3724452976.000003 s since 1904-01-01), "数值 2"=-40.9000015258789}, {"数值"=timestamp(3724453076.000003 s since 1904-01-01), "数值 2"=-40.0999984741211}, {"数值"=timestamp(3724453176.000003 s since 1904-01-01), "数值 2"=-38.0}, {"数值"=timestamp(3724453276.000003 s since 1904-01-01), "数值 2"=-38.0999984741211}, {"数值"=timestamp(3724453376.000003 s since 1904-01-01), "数值 2"=-39.4000015258789}, {"数值"=timestamp(3724453476.000003 s since 1904-01-01), "数值 2"=-40.5}, {"数值"=timestamp(3724453576.000003 s since 1904-01-01), "数值 2"=-40.9000015258789}, {"数值"=timestamp(3724453676.000003 s since 1904-01-01), "数值 2"=-40.7000007629395}, {"数值"=timestamp(3724453776.000003 s since 1904-01-01), "数值 2"=-39.2999992370605}, {"数值"=timestamp(3724453876.000003 s since 1904-01-01), "数值 2"=-38.7999992370605}, {"数值"=timestamp(3724453976.000003 s since 1904-01-01), "数值 2"=-40.2000007629395}, {"数值"=timestamp(3724454076.000003 s since 1904-01-01), "数值 2"=-41.0999984741211}, {"数值"=timestamp(3724454176.000003 s since 1904-01-01), "数值 2"=-41.2999992370605}, {"数值"=timestamp(3724454276.000003 s since 1904-01-01), "数值 2"=-40.0}, {"数值"=timestamp(3724454376.000003 s since 1904-01-01), "数值 2"=-38.5999984741211}, {"数值"=timestamp(3724454476.000003 s since 1904-01-01), "数值 2"=-38.5999984741211}, {"数值"=timestamp(3724454576.000003 s since 1904-01-01), "数值 2"=-40.5999984741211}, {"数值"=timestamp(3724454676.000003 s since 1904-01-01), "数值 2"=-41.0999984741211}, {"数值"=timestamp(3724454776.000003 s since 1904-01-01), "数值 2"=-40.7999992370605}, {"数值"=timestamp(3724454876.000003 s since 1904-01-01), "数值 2"=-39.0}, {"数值"=timestamp(3724454976.000003 s since 1904-01-01), "数值 2"=-38.7000007629395}, {"数值"=timestamp(3724455076.000003 s since 1904-01-01), "数值 2"=-39.7999992370605}, {"数值"=timestamp(3724455176.000003 s since 1904-01-01), "数值 2"=-41.0}, {"数值"=timestamp(3724455276.000003 s since 1904-01-01), "数值 2"=-41.0999984741211}, {"数值"=timestamp(3724455376.000003 s since 1904-01-01), "数值 2"=-40.2000007629395}, {"数值"=timestamp(3724455476.000003 s since 1904-01-01), "数值 2"=65.0}, {"数值"=timestamp(3724455576.000003 s since 1904-01-01), "数值 2"=86.3000030517578}, {"数值"=timestamp(3724455676.000003 s since 1904-01-01), "数值 2"=85.1999969482422}, {"数值"=timestamp(3724455776.000003 s since 1904-01-01), "数值 2"=85.1999969482422}, {"数值"=timestamp(3724455876.000003 s since 1904-01-01), "数值 2"=85.0}, {"数值"=timestamp(3724455976.000003 s since 1904-01-01), "数值 2"=85.0999984741211}, {"数值"=timestamp(3724456076.000003 s since 1904-01-01), "数值 2"=85.0}, {"数值"=timestamp(3724456176.000003 s since 1904-01-01), "数值 2"=85.0}, {"数值"=timestamp(3724456276.000003 s since 1904-01-01), "数值 2"=85.0}, {"数值"=timestamp(3724456376.000003 s since 1904-01-01), "数值 2"=85.0}, {"数值"=timestamp(3724456476.000003 s since 1904-01-01), "数值 2"=85.0}, {"数值"=timestamp(3724456576.000003 s since 1904-01-01), "数值 2"=85.0}, {"数值"=timestamp(3724456676.000003 s since 1904-01-01), "数值 2"=85.0}, {"数值"=timestamp(3724456776.000003 s since 1904-01-01), "数值 2"=85.0999984741211}, {"数值"=timestamp(3724456876.000003 s since 1904-01-01), "数值 2"=85.0}, {"数值"=timestamp(3724456976.000003 s since 1904-01-01), "数值 2"=84.9000015258789}, {"数值"=timestamp(3724457076.000003 s since 1904-01-01), "数值 2"=84.9000015258789}, {"数值"=timestamp(3724457176.000003 s since 1904-01-01), "数值 2"=85.0}, {"数值"=timestamp(3724457276.000003 s since 1904-01-01), "数值 2"=-11.1999998092651}, {"数值"=timestamp(3724457376.000003 s since 1904-01-01), "数值 2"=-42.9000015258789}, {"数值"=timestamp(3724457476.000003 s since 1904-01-01), "数值 2"=-40.9000015258789}, {"数值"=timestamp(3724457576.000003 s since 1904-01-01), "数值 2"=-39.7999992370605}, {"数值"=timestamp(3724457676.000003 s since 1904-01-01), "数值 2"=-38.0}, {"数值"=timestamp(3724457776.000003 s since 1904-01-01), "数值 2"=-38.2000007629395}, {"数值"=timestamp(3724457876.000003 s since 1904-01-01), "数值 2"=-39.5999984741211}, {"数值"=timestamp(3724457976.000003 s since 1904-01-01), "数值 2"=-40.5}, {"数值"=timestamp(3724458076.000003 s since 1904-01-01), "数值 2"=-40.7999992370605}, {"数值"=timestamp(3724458176.000003 s since 1904-01-01), "数值 2"=-40.5999984741211}, {"数值"=timestamp(3724458276.000003 s since 1904-01-01), "数值 2"=-39.4000015258789}, {"数值"=timestamp(3724458376.000003 s since 1904-01-01), "数值 2"=-38.9000015258789}, {"数值"=timestamp(3724458476.000003 s since 1904-01-01), "数值 2"=-40.2000007629395}, {"数值"=timestamp(3724458576.000003 s since 1904-01-01), "数值 2"=-41.0}, {"数值"=timestamp(3724458676.000003 s since 1904-01-01), "数值 2"=-41.2000007629395}, {"数值"=timestamp(3724458776.000003 s since 1904-01-01), "数值 2"=-39.9000015258789}, {"数值"=timestamp(3724458876.000003 s since 1904-01-01), "数值 2"=-38.7000007629395}, {"数值"=timestamp(3724458976.000003 s since 1904-01-01), "数值 2"=-39.0}, {"数值"=timestamp(3724459076.000003 s since 1904-01-01), "数值 2"=-40.7999992370605}, {"数值"=timestamp(3724459176.000003 s since 1904-01-01), "数值 2"=-41.0999984741211}, {"数值"=timestamp(3724459276.000003 s since 1904-01-01), "数值 2"=-40.5999984741211}, {"数值"=timestamp(3724459376.000003 s since 1904-01-01), "数值 2"=-38.7000007629395}, {"数值"=timestamp(3724459476.000003 s since 1904-01-01), "数值 2"=-38.7000007629395}, {"数值"=timestamp(3724459576.000003 s since 1904-01-01), "数值 2"=-40.0}, {"数值"=timestamp(3724459676.000003 s since 1904-01-01), "数值 2"=-41.0999984741211}, {"数值"=timestamp(3724459776.000003 s since 1904-01-01), "数值 2"=-40.7999992370605}, {"数值"=timestamp(3724459876.000003 s since 1904-01-01), "数值 2"=-39.7000007629395}, {"数值"=timestamp(3724459976.000003 s since 1904-01-01), "数值 2"=79.5999984741211}, {"数值"=timestamp(3724460076.000003 s since 1904-01-01), "数值 2"=86.0999984741211}, {"数值"=timestamp(3724460176.000003 s since 1904-01-01), "数值 2"=85.3000030517578}, {"数值"=timestamp(3724460276.000003 s since 1904-01-01), "数值 2"=85.0999984741211}, {"数值"=timestamp(3724460376.000003 s since 1904-01-01), "数值 2"=84.9000015258789}, {"数值"=timestamp(3724460476.000003 s since 1904-01-01), "数值 2"=84.9000015258789}, {"数值"=timestamp(3724460576.000003 s since 1904-01-01), "数值 2"=85.0}, {"数值"=timestamp(3724460676.000003 s since 1904-01-01), "数值 2"=85.0}, {"数值"=timestamp(3724460776.000003 s since 1904-01-01), "数值 2"=85.0}, {"数值"=timestamp(3724460876.000003 s since 1904-01-01), "数值 2"=85.0}, {"数值"=timestamp(3724460976.000003 s since 1904-01-01), "数值 2"=85.0}, {"数值"=timestamp(3724461076.000003 s since 1904-01-01), "数值 2"=85.0}, {"数值"=timestamp(3724461176.000003 s since 1904-01-01), "数值 2"=85.0}, {"数值"=timestamp(3724461276.000003 s since 1904-01-01), "数值 2"=84.9000015258789}, {"数值"=timestamp(3724461376.000003 s since 1904-01-01), "数值 2"=85.0}, {"数值"=timestamp(3724461476.000003 s since 1904-01-01), "数值 2"=84.9000015258789}, {"数值"=timestamp(3724461576.000003 s since 1904-01-01), "数值 2"=85.0}, {"数值"=timestamp(3724461676.000003 s since 1904-01-01), "数值 2"=85.0}, {"数值"=timestamp(3724461776.000003 s since 1904-01-01), "数值 2"=60.2000007629395}, {"数值"=timestamp(3724461876.000003 s since 1904-01-01), "数值 2"=-42.5}, {"数值"=timestamp(3724461976.000003 s since 1904-01-01), "数值 2"=-40.7000007629395}, {"数值"=timestamp(3724462076.000003 s since 1904-01-01), "数值 2"=-40.2000007629395}, {"数值"=timestamp(3724462176.000003 s since 1904-01-01), "数值 2"=-38.0}, {"数值"=timestamp(3724462276.000003 s since 1904-01-01), "数值 2"=-38.4000015258789}, {"数值"=timestamp(3724462376.000003 s since 1904-01-01), "数值 2"=-39.0999984741211}, {"数值"=timestamp(3724462476.000003 s since 1904-01-01), "数值 2"=-40.7999992370605}, {"数值"=timestamp(3724462576.000003 s since 1904-01-01), "数值 2"=-41.2000007629395}, {"数值"=timestamp(3724462676.000003 s since 1904-01-01), "数值 2"=-40.7000007629395}, {"数值"=timestamp(3724462776.000003 s since 1904-01-01), "数值 2"=-38.9000015258789}, {"数值"=timestamp(3724462876.000003 s since 1904-01-01), "数值 2"=-38.7000007629395}, {"数值"=timestamp(3724462976.000003 s since 1904-01-01), "数值 2"=-40.0999984741211}, {"数值"=timestamp(3724463076.000003 s since 1904-01-01), "数值 2"=-41.0999984741211}, {"数值"=timestamp(3724463176.000003 s since 1904-01-01), "数值 2"=-40.9000015258789}, {"数值"=timestamp(3724463276.000003 s since 1904-01-01), "数值 2"=-39.9000015258789}, {"数值"=timestamp(3724463376.000003 s since 1904-01-01), "数值 2"=-38.5999984741211}, {"数值"=timestamp(3724463476.000003 s since 1904-01-01), "数值 2"=-39.5999984741211}, {"数值"=timestamp(3724463576.000003 s since 1904-01-01), "数值 2"=-40.9000015258789}, {"数值"=timestamp(3724463676.000003 s since 1904-01-01), "数值 2"=-41.0}, {"数值"=timestamp(3724463776.000003 s since 1904-01-01), "数值 2"=-40.2000007629395}, {"数值"=timestamp(3724463876.000003 s since 1904-01-01), "数值 2"=-38.7999992370605}, {"数值"=timestamp(3724463976.000003 s since 1904-01-01), "数值 2"=-39.0}, {"数值"=timestamp(3724464076.000003 s since 1904-01-01), "数值 2"=-40.5}, {"数值"=timestamp(3724464176.000003 s since 1904-01-01), "数值 2"=-40.9000015258789}, {"数值"=timestamp(3724464276.000003 s since 1904-01-01), "数值 2"=-40.5999984741211}, {"数值"=timestamp(3724464376.000003 s since 1904-01-01), "数值 2"=-39.0999984741211}, {"数值"=timestamp(3724464476.000003 s since 1904-01-01), "数值 2"=11.3999996185303}, {"数值"=timestamp(3724464576.000003 s since 1904-01-01), "数值 2"=86.0}, {"数值"=timestamp(3724464676.000003 s since 1904-01-01), "数值 2"=85.1999969482422}, {"数值"=timestamp(3724464776.000003 s since 1904-01-01), "数值 2"=85.1999969482422}, {"数值"=timestamp(3724464876.000003 s since 1904-01-01), "数值 2"=85.0}, {"数值"=timestamp(3724464976.000003 s since 1904-01-01), "数值 2"=85.0}, {"数值"=timestamp(3724465076.000003 s since 1904-01-01), "数值 2"=85.0}, {"数值"=timestamp(3724465176.000003 s since 1904-01-01), "数值 2"=85.0}, {"数值"=timestamp(3724465276.000003 s since 1904-01-01), "数值 2"=85.0}, {"数值"=timestamp(3724465376.000003 s since 1904-01-01), "数值 2"=85.0}, {"数值"=timestamp(3724465476.000003 s since 1904-01-01), "数值 2"=85.0}, {"数值"=timestamp(3724465576.000003 s since 1904-01-01), "数值 2"=85.0}, {"数值"=timestamp(3724465676.000003 s since 1904-01-01), "数值 2"=85.0}, {"数值"=timestamp(3724465776.000003 s since 1904-01-01), "数值 2"=85.0}, {"数值"=timestamp(3724465876.000003 s since 1904-01-01), "数值 2"=85.0}, {"数值"=timestamp(3724465976.000003 s since 1904-01-01), "数值 2"=85.0999984741211}, {"数值"=timestamp(3724466076.000003 s since 1904-01-01), "数值 2"=84.9000015258789}, {"数值"=timestamp(3724466176.000003 s since 1904-01-01), "数值 2"=85.0}, {"数值"=timestamp(3724466276.000003 s since 1904-01-01), "数值 2"=27.6000003814697}, {"数值"=timestamp(3724466376.000003 s since 1904-01-01), "数值 2"=-42.0999984741211}, {"数值"=timestamp(3724466476.000003 s since 1904-01-01), "数值 2"=-40.7999992370605}, {"数值"=timestamp(3724466576.000003 s since 1904-01-01), "数值 2"=-40.2000007629395}, {"数值"=timestamp(3724466676.000003 s since 1904-01-01), "数值 2"=-38.0}, {"数值"=timestamp(3724466776.000003 s since 1904-01-01), "数值 2"=-38.5999984741211}, {"数值"=timestamp(3724466876.000003 s since 1904-01-01), "数值 2"=-39.2999992370605}, {"数值"=timestamp(3724466976.000003 s since 1904-01-01), "数值 2"=-40.9000015258789}, {"数值"=timestamp(3724467076.000003 s since 1904-01-01), "数值 2"=-41.2999992370605}, {"数值"=timestamp(3724467176.000003 s since 1904-01-01), "数值 2"=-40.7999992370605}, {"数值"=timestamp(3724467276.000003 s since 1904-01-01), "数值 2"=-39.4000015258789}, {"数值"=timestamp(3724467376.000003 s since 1904-01-01), "数值 2"=-38.7000007629395}, {"数值"=timestamp(3724467476.000003 s since 1904-01-01), "数值 2"=-39.7000007629395}, {"数值"=timestamp(3724467576.000003 s since 1904-01-01), "数值 2"=-41.0}, {"数值"=timestamp(3724467676.000003 s since 1904-01-01), "数值 2"=-41.0999984741211}, {"数值"=timestamp(3724467776.000003 s since 1904-01-01), "数值 2"=-40.2000007629395}, {"数值"=timestamp(3724467876.000003 s since 1904-01-01), "数值 2"=-38.7999992370605}, {"数值"=timestamp(3724467976.000003 s since 1904-01-01), "数值 2"=-38.9000015258789}, {"数值"=timestamp(3724468076.000003 s since 1904-01-01), "数值 2"=-40.2999992370605}, {"数值"=timestamp(3724468176.000003 s since 1904-01-01), "数值 2"=-41.2000007629395}, {"数值"=timestamp(3724468276.000003 s since 1904-01-01), "数值 2"=-40.9000015258789}, {"数值"=timestamp(3724468376.000003 s since 1904-01-01), "数值 2"=-39.7000007629395}, {"数值"=timestamp(3724468476.000003 s since 1904-01-01), "数值 2"=-38.5999984741211}, {"数值"=timestamp(3724468576.000003 s since 1904-01-01), "数值 2"=-39.4000015258789}, {"数值"=timestamp(3724468676.000003 s since 1904-01-01), "数值 2"=-40.9000015258789}, {"数值"=timestamp(3724468776.000003 s since 1904-01-01), "数值 2"=-41.4000015258789}, {"数值"=timestamp(3724468876.000003 s since 1904-01-01), "数值 2"=-40.4000015258789}, {"数值"=timestamp(3724468976.000003 s since 1904-01-01), "数值 2"=45.0999984741211}, {"数值"=timestamp(3724469076.000003 s since 1904-01-01), "数值 2"=86.4000015258789}, {"数值"=timestamp(3724469176.000003 s since 1904-01-01), "数值 2"=85.1999969482422}, {"数值"=timestamp(3724469276.000003 s since 1904-01-01), "数值 2"=85.0}, {"数值"=timestamp(3724469376.000003 s since 1904-01-01), "数值 2"=85.0999984741211}, {"数值"=timestamp(3724469476.000003 s since 1904-01-01), "数值 2"=85.0}, {"数值"=timestamp(3724469576.000003 s since 1904-01-01), "数值 2"=85.0}, {"数值"=timestamp(3724469676.000003 s since 1904-01-01), "数值 2"=85.0}, {"数值"=timestamp(3724469776.000003 s since 1904-01-01), "数值 2"=85.0}, {"数值"=timestamp(3724469876.000003 s since 1904-01-01), "数值 2"=85.0999984741211}, {"数值"=timestamp(3724469976.000003 s since 1904-01-01), "数值 2"=85.0999984741211}, {"数值"=timestamp(3724470076.000003 s since 1904-01-01), "数值 2"=85.0}, {"数值"=timestamp(3724470176.000003 s since 1904-01-01), "数值 2"=85.0}, {"数值"=timestamp(3724470276.000003 s since 1904-01-01), "数值 2"=84.9000015258789}, {"数值"=timestamp(3724470376.000003 s since 1904-01-01), "数值 2"=85.0}, {"数值"=timestamp(3724470476.000003 s since 1904-01-01), "数值 2"=85.0}, {"数值"=timestamp(3724470576.000003 s since 1904-01-01), "数值 2"=85.0}, {"数值"=timestamp(3724470676.000003 s since 1904-01-01), "数值 2"=85.0999984741211}, {"数值"=timestamp(3724470776.000003 s since 1904-01-01), "数值 2"=8.0}, {"数值"=timestamp(3724470876.000003 s since 1904-01-01), "数值 2"=-43.0}, {"数值"=timestamp(3724470976.000003 s since 1904-01-01), "数值 2"=-40.7999992370605}, {"数值"=timestamp(3724471076.000003 s since 1904-01-01), "数值 2"=-40.4000015258789}, {"数值"=timestamp(3724471176.000003 s since 1904-01-01), "数值 2"=-38.0}, {"数值"=timestamp(3724471276.000003 s since 1904-01-01), "数值 2"=-38.4000015258789}, {"数值"=timestamp(3724471376.000003 s since 1904-01-01), "数值 2"=-39.2000007629395}, {"数值"=timestamp(3724471476.000003 s since 1904-01-01), "数值 2"=-40.7999992370605}, {"数值"=timestamp(3724471576.000003 s since 1904-01-01), "数值 2"=-41.0999984741211}, {"数值"=timestamp(3724471676.000003 s since 1904-01-01), "数值 2"=-40.5999984741211}, {"数值"=timestamp(3724471776.000003 s since 1904-01-01), "数值 2"=-39.0999984741211}, {"数值"=timestamp(3724471876.000003 s since 1904-01-01), "数值 2"=-39.0}, {"数值"=timestamp(3724471976.000003 s since 1904-01-01), "数值 2"=-40.2000007629395}, {"数值"=timestamp(3724472076.000003 s since 1904-01-01), "数值 2"=-40.9000015258789}, {"数值"=timestamp(3724472176.000003 s since 1904-01-01), "数值 2"=-40.7999992370605}, {"数值"=timestamp(3724472276.000003 s since 1904-01-01), "数值 2"=-39.7000007629395}, {"数值"=timestamp(3724472376.000003 s since 1904-01-01), "数值 2"=-38.5999984741211}, {"数值"=timestamp(3724472476.000003 s since 1904-01-01), "数值 2"=-39.7999992370605}, {"数值"=timestamp(3724472576.000003 s since 1904-01-01), "数值 2"=-40.9000015258789}, {"数值"=timestamp(3724472676.000003 s since 1904-01-01), "数值 2"=-41.2000007629395}, {"数值"=timestamp(3724472776.000003 s since 1904-01-01), "数值 2"=-40.2000007629395}, {"数值"=timestamp(3724472876.000003 s since 1904-01-01), "数值 2"=-38.5999984741211}, {"数值"=timestamp(3724472976.000003 s since 1904-01-01), "数值 2"=-38.9000015258789}, {"数值"=timestamp(3724473076.000003 s since 1904-01-01), "数值 2"=-40.5999984741211}, {"数值"=timestamp(3724473176.000003 s since 1904-01-01), "数值 2"=-41.2999992370605}, {"数值"=timestamp(3724473276.000003 s since 1904-01-01), "数值 2"=-40.9000015258789}, {"数值"=timestamp(3724473376.000003 s since 1904-01-01), "数值 2"=-39.2000007629395}, {"数值"=timestamp(3724473476.000003 s since 1904-01-01), "数值 2"=65.8000030517578}, {"数值"=timestamp(3724473576.000003 s since 1904-01-01), "数值 2"=86.4000015258789}, {"数值"=timestamp(3724473676.000003 s since 1904-01-01), "数值 2"=85.1999969482422}, {"数值"=timestamp(3724473776.000003 s since 1904-01-01), "数值 2"=85.0999984741211}, {"数值"=timestamp(3724473876.000003 s since 1904-01-01), "数值 2"=84.9000015258789}, {"数值"=timestamp(3724473976.000003 s since 1904-01-01), "数值 2"=84.9000015258789}, {"数值"=timestamp(3724474076.000003 s since 1904-01-01), "数值 2"=85.0}, {"数值"=timestamp(3724474176.000003 s since 1904-01-01), "数值 2"=85.0}, {"数值"=timestamp(3724474276.000003 s since 1904-01-01), "数值 2"=85.0}, {"数值"=timestamp(3724474376.000003 s since 1904-01-01), "数值 2"=85.0}, {"数值"=timestamp(3724474476.000003 s since 1904-01-01), "数值 2"=85.0}, {"数值"=timestamp(3724474576.000003 s since 1904-01-01), "数值 2"=85.0999984741211}, {"数值"=timestamp(3724474676.000003 s since 1904-01-01), "数值 2"=85.0}, {"数值"=timestamp(3724474776.000003 s since 1904-01-01), "数值 2"=85.0}, {"数值"=timestamp(3724474876.000003 s since 1904-01-01), "数值 2"=85.0}, {"数值"=timestamp(3724474976.000003 s since 1904-01-01), "数值 2"=85.0999984741211}, {"数值"=timestamp(3724475076.000003 s since 1904-01-01), "数值 2"=85.0}, {"数值"=timestamp(3724475176.000003 s since 1904-01-01), "数值 2"=85.0}, {"数值"=timestamp(3724475276.000003 s since 1904-01-01), "数值 2"=-8.80000019073486}, {"数值"=timestamp(3724475376.000003 s since 1904-01-01), "数值 2"=-43.7000007629395}, {"数值"=timestamp(3724475476.000003 s since 1904-01-01), "数值 2"=-41.2999992370605}, {"数值"=timestamp(3724475576.000003 s since 1904-01-01), "数值 2"=-40.4000015258789}, {"数值"=timestamp(3724475676.000003 s since 1904-01-01), "数值 2"=-38.0}, {"数值"=timestamp(3724475776.000003 s since 1904-01-01), "数值 2"=-38.5}, {"数值"=timestamp(3724475876.000003 s since 1904-01-01), "数值 2"=-39.2999992370605}, {"数值"=timestamp(3724475976.000003 s since 1904-01-01), "数值 2"=-40.4000015258789}, {"数值"=timestamp(3724476076.000003 s since 1904-01-01), "数值 2"=-41.2999992370605}, {"数值"=timestamp(3724476176.000003 s since 1904-01-01), "数值 2"=-40.9000015258789}, {"数值"=timestamp(3724476276.000003 s since 1904-01-01), "数值 2"=-39.7999992370605}, {"数值"=timestamp(3724476376.000003 s since 1904-01-01), "数值 2"=-38.5}, {"数值"=timestamp(3724476476.000003 s since 1904-01-01), "数值 2"=-39.5999984741211}, {"数值"=timestamp(3724476576.000003 s since 1904-01-01), "数值 2"=-40.7999992370605}, {"数值"=timestamp(3724476676.000003 s since 1904-01-01), "数值 2"=-41.0999984741211}, {"数值"=timestamp(3724476776.000003 s since 1904-01-01), "数值 2"=-40.2999992370605}, {"数值"=timestamp(3724476876.000003 s since 1904-01-01), "数值 2"=-38.7000007629395}, {"数值"=timestamp(3724476976.000003 s since 1904-01-01), "数值 2"=-38.7999992370605}, {"数值"=timestamp(3724477076.000003 s since 1904-01-01), "数值 2"=-40.7000007629395}, {"数值"=timestamp(3724477176.000003 s since 1904-01-01), "数值 2"=-41.0999984741211}, {"数值"=timestamp(3724477276.000003 s since 1904-01-01), "数值 2"=-40.7000007629395}, {"数值"=timestamp(3724477376.000003 s since 1904-01-01), "数值 2"=-39.0}, {"数值"=timestamp(3724477476.000003 s since 1904-01-01), "数值 2"=-38.7000007629395}, {"数值"=timestamp(3724477576.000003 s since 1904-01-01), "数值 2"=-39.7999992370605}, {"数值"=timestamp(3724477676.000003 s since 1904-01-01), "数值 2"=-41.0999984741211}, {"数值"=timestamp(3724477776.000003 s since 1904-01-01), "数值 2"=-41.0999984741211}, {"数值"=timestamp(3724477876.000003 s since 1904-01-01), "数值 2"=-40.0}, {"数值"=timestamp(3724477976.000003 s since 1904-01-01), "数值 2"=77.5}, {"数值"=timestamp(3724478076.000003 s since 1904-01-01), "数值 2"=86.1999969482422}, {"数值"=timestamp(3724478176.000003 s since 1904-01-01), "数值 2"=85.1999969482422}, {"数值"=timestamp(3724478276.000003 s since 1904-01-01), "数值 2"=85.0999984741211}, {"数值"=timestamp(3724478376.000003 s since 1904-01-01), "数值 2"=85.0}, {"数值"=timestamp(3724478476.000003 s since 1904-01-01), "数值 2"=85.0}, {"数值"=timestamp(3724478576.000003 s since 1904-01-01), "数值 2"=85.0}, {"数值"=timestamp(3724478676.000003 s since 1904-01-01), "数值 2"=85.0}, {"数值"=timestamp(3724478776.000003 s since 1904-01-01), "数值 2"=85.0}, {"数值"=timestamp(3724478876.000003 s since 1904-01-01), "数值 2"=85.0}, {"数值"=timestamp(3724478976.000003 s since 1904-01-01), "数值 2"=85.0}, {"数值"=timestamp(3724479076.000003 s since 1904-01-01), "数值 2"=85.0}, {"数值"=timestamp(3724479176.000003 s since 1904-01-01), "数值 2"=85.0}, {"数值"=timestamp(3724479276.000003 s since 1904-01-01), "数值 2"=85.0}, {"数值"=timestamp(3724479376.000003 s since 1904-01-01), "数值 2"=85.0}, {"数值"=timestamp(3724479476.000003 s since 1904-01-01), "数值 2"=84.9000015258789}, {"数值"=timestamp(3724479576.000003 s since 1904-01-01), "数值 2"=84.9000015258789}, {"数值"=timestamp(3724479676.000003 s since 1904-01-01), "数值 2"=85.0}, {"数值"=timestamp(3724479776.000003 s since 1904-01-01), "数值 2"=-21.0}, {"数值"=timestamp(3724479876.000003 s since 1904-01-01), "数值 2"=-42.5999984741211}, {"数值"=timestamp(3724479976.000003 s since 1904-01-01), "数值 2"=-40.5999984741211}, {"数值"=timestamp(3724480076.000003 s since 1904-01-01), "数值 2"=-39.9000015258789}, {"数值"=timestamp(3724480176.000003 s since 1904-01-01), "数值 2"=-37.9000015258789}, {"数值"=timestamp(3724480276.000003 s since 1904-01-01), "数值 2"=-38.4000015258789}, {"数值"=timestamp(3724480376.000003 s since 1904-01-01), "数值 2"=-39.5}, {"数值"=timestamp(3724480476.000003 s since 1904-01-01), "数值 2"=-40.7999992370605}, {"数值"=timestamp(3724480576.000003 s since 1904-01-01), "数值 2"=-41.0999984741211}, {"数值"=timestamp(3724480676.000003 s since 1904-01-01), "数值 2"=-40.2999992370605}, {"数值"=timestamp(3724480776.000003 s since 1904-01-01), "数值 2"=-39.0}, {"数值"=timestamp(3724480876.000003 s since 1904-01-01), "数值 2"=-39.2000007629395}, {"数值"=timestamp(3724480976.000003 s since 1904-01-01), "数值 2"=-39.9000015258789}, {"数值"=timestamp(3724481076.000003 s since 1904-01-01), "数值 2"=-40.9000015258789}, {"数值"=timestamp(3724481176.000003 s since 1904-01-01), "数值 2"=-41.2000007629395}, {"数值"=timestamp(3724481276.000003 s since 1904-01-01), "数值 2"=-40.0}, {"数值"=timestamp(3724481376.000003 s since 1904-01-01), "数值 2"=-38.5999984741211}, {"数值"=timestamp(3724481476.000003 s since 1904-01-01), "数值 2"=-38.7999992370605}, {"数值"=timestamp(3724481576.000003 s since 1904-01-01), "数值 2"=-40.5}, {"数值"=timestamp(3724481676.000003 s since 1904-01-01), "数值 2"=-41.0999984741211}, {"数值"=timestamp(3724481776.000003 s since 1904-01-01), "数值 2"=-40.7000007629395}, {"数值"=timestamp(3724481876.000003 s since 1904-01-01), "数值 2"=-39.4000015258789}, {"数值"=timestamp(3724481976.000003 s since 1904-01-01), "数值 2"=-38.7000007629395}, {"数值"=timestamp(3724482076.000003 s since 1904-01-01), "数值 2"=-40.0}, {"数值"=timestamp(3724482176.000003 s since 1904-01-01), "数值 2"=-40.9000015258789}, {"数值"=timestamp(3724482276.000003 s since 1904-01-01), "数值 2"=-40.9000015258789}, {"数值"=timestamp(3724482376.000003 s since 1904-01-01), "数值 2"=-39.7999992370605}, {"数值"=timestamp(3724482476.000003 s since 1904-01-01), "数值 2"=11.6999998092651}, {"数值"=timestamp(3724482576.000003 s since 1904-01-01), "数值 2"=86.0}, {"数值"=timestamp(3724482676.000003 s since 1904-01-01), "数值 2"=85.1999969482422}, {"数值"=timestamp(3724482776.000003 s since 1904-01-01), "数值 2"=85.0999984741211}, {"数值"=timestamp(3724482876.000003 s since 1904-01-01), "数值 2"=84.9000015258789}, {"数值"=timestamp(3724482976.000003 s since 1904-01-01), "数值 2"=84.9000015258789}, {"数值"=timestamp(3724483076.000003 s since 1904-01-01), "数值 2"=85.0}, {"数值"=timestamp(3724483176.000003 s since 1904-01-01), "数值 2"=85.0}, {"数值"=timestamp(3724483276.000003 s since 1904-01-01), "数值 2"=85.0}, {"数值"=timestamp(3724483376.000003 s since 1904-01-01), "数值 2"=85.0}, {"数值"=timestamp(3724483476.000003 s since 1904-01-01), "数值 2"=85.0}, {"数值"=timestamp(3724483576.000003 s since 1904-01-01), "数值 2"=85.0}, {"数值"=timestamp(3724483676.000003 s since 1904-01-01), "数值 2"=85.0}, {"数值"=timestamp(3724483776.000003 s since 1904-01-01), "数值 2"=85.0}, {"数值"=timestamp(3724483876.000003 s since 1904-01-01), "数值 2"=85.0}, {"数值"=timestamp(3724483976.000003 s since 1904-01-01), "数值 2"=85.0}, {"数值"=timestamp(3724484076.000003 s since 1904-01-01), "数值 2"=84.9000015258789}, {"数值"=timestamp(3724484176.000003 s since 1904-01-01), "数值 2"=84.9000015258789}, {"数值"=timestamp(3724484276.000003 s since 1904-01-01), "数值 2"=31.2999992370605}, {"数值"=timestamp(3724484376.000003 s since 1904-01-01), "数值 2"=-42.0}, {"数值"=timestamp(3724484476.000003 s since 1904-01-01), "数值 2"=-40.7000007629395}, {"数值"=timestamp(3724484576.000003 s since 1904-01-01), "数值 2"=-40.2000007629395}, {"数值"=timestamp(3724484676.000003 s since 1904-01-01), "数值 2"=-38.0}, {"数值"=timestamp(3724484776.000003 s since 1904-01-01), "数值 2"=-38.2000007629395}, {"数值"=timestamp(3724484876.000003 s since 1904-01-01), "数值 2"=-38.9000015258789}, {"数值"=timestamp(3724484976.000003 s since 1904-01-01), "数值 2"=-40.7000007629395}, {"数值"=timestamp(3724485076.000003 s since 1904-01-01), "数值 2"=-41.0999984741211}, {"数值"=timestamp(3724485176.000003 s since 1904-01-01), "数值 2"=-40.7000007629395}, {"数值"=timestamp(3724485276.000003 s since 1904-01-01), "数值 2"=-38.9000015258789}, {"数值"=timestamp(3724485376.000003 s since 1904-01-01), "数值 2"=-38.7999992370605}, {"数值"=timestamp(3724485476.000003 s since 1904-01-01), "数值 2"=-40.4000015258789}, {"数值"=timestamp(3724485576.000003 s since 1904-01-01), "数值 2"=-41.0999984741211}, {"数值"=timestamp(3724485676.000003 s since 1904-01-01), "数值 2"=-40.7999992370605}, {"数值"=timestamp(3724485776.000003 s since 1904-01-01), "数值 2"=-39.5999984741211}, {"数值"=timestamp(3724485876.000003 s since 1904-01-01), "数值 2"=-38.7000007629395}, {"数值"=timestamp(3724485976.000003 s since 1904-01-01), "数值 2"=-39.7000007629395}, {"数值"=timestamp(3724486076.000003 s since 1904-01-01), "数值 2"=-40.7999992370605}, {"数值"=timestamp(3724486176.000003 s since 1904-01-01), "数值 2"=-41.2999992370605}, {"数值"=timestamp(3724486276.000003 s since 1904-01-01), "数值 2"=-40.4000015258789}, {"数值"=timestamp(3724486376.000003 s since 1904-01-01), "数值 2"=-39.0}, {"数值"=timestamp(3724486476.000003 s since 1904-01-01), "数值 2"=-38.7999992370605}, {"数值"=timestamp(3724486576.000003 s since 1904-01-01), "数值 2"=-40.4000015258789}, {"数值"=timestamp(3724486676.000003 s since 1904-01-01), "数值 2"=-41.2000007629395}, {"数值"=timestamp(3724486776.000003 s since 1904-01-01), "数值 2"=-41.0}, {"数值"=timestamp(3724486876.000003 s since 1904-01-01), "数值 2"=-40.0}, {"数值"=timestamp(3724486976.000003 s since 1904-01-01), "数值 2"=43.7000007629395}, {"数值"=timestamp(3724487076.000003 s since 1904-01-01), "数值 2"=85.6999969482422}, {"数值"=timestamp(3724487176.000003 s since 1904-01-01), "数值 2"=85.1999969482422}, {"数值"=timestamp(3724487276.000003 s since 1904-01-01), "数值 2"=85.0999984741211}, {"数值"=timestamp(3724487376.000003 s since 1904-01-01), "数值 2"=84.9000015258789}, {"数值"=timestamp(3724487476.000003 s since 1904-01-01), "数值 2"=84.9000015258789}, {"数值"=timestamp(3724487576.000003 s since 1904-01-01), "数值 2"=85.0}, {"数值"=timestamp(3724487676.000003 s since 1904-01-01), "数值 2"=85.0}, {"数值"=timestamp(3724487776.000003 s since 1904-01-01), "数值 2"=85.0}, {"数值"=timestamp(3724487876.000003 s since 1904-01-01), "数值 2"=85.0}, {"数值"=timestamp(3724487976.000003 s since 1904-01-01), "数值 2"=85.0}, {"数值"=timestamp(3724488076.000003 s since 1904-01-01), "数值 2"=85.0}, {"数值"=timestamp(3724488176.000003 s since 1904-01-01), "数值 2"=84.9000015258789}, {"数值"=timestamp(3724488276.000003 s since 1904-01-01), "数值 2"=85.0}, {"数值"=timestamp(3724488376.000003 s since 1904-01-01), "数值 2"=85.0}, {"数值"=timestamp(3724488476.000003 s since 1904-01-01), "数值 2"=85.0}, {"数值"=timestamp(3724488576.000003 s since 1904-01-01), "数值 2"=85.0999984741211}, {"数值"=timestamp(3724488676.000003 s since 1904-01-01), "数值 2"=85.0}, {"数值"=timestamp(3724488776.000003 s since 1904-01-01), "数值 2"=7.19999980926514}, {"数值"=timestamp(3724488876.000003 s since 1904-01-01), "数值 2"=-43.2000007629395}, {"数值"=timestamp(3724488976.000003 s since 1904-01-01), "数值 2"=-40.4000015258789}, {"数值"=timestamp(3724489076.000003 s since 1904-01-01), "数值 2"=-40.2999992370605}, {"数值"=timestamp(3724489176.000003 s since 1904-01-01), "数值 2"=-38.0}, {"数值"=timestamp(3724489276.000003 s since 1904-01-01), "数值 2"=-38.4000015258789}, {"数值"=timestamp(3724489376.000003 s since 1904-01-01), "数值 2"=-39.2000007629395}, {"数值"=timestamp(3724489476.000003 s since 1904-01-01), "数值 2"=-40.5}, {"数值"=timestamp(3724489576.000003 s since 1904-01-01), "数值 2"=-41.2000007629395}, {"数值"=timestamp(3724489676.000003 s since 1904-01-01), "数值 2"=-40.7999992370605}, {"数值"=timestamp(3724489776.000003 s since 1904-01-01), "数值 2"=-39.5}, {"数值"=timestamp(3724489876.000003 s since 1904-01-01), "数值 2"=-38.5999984741211}, {"数值"=timestamp(3724489976.000003 s since 1904-01-01), "数值 2"=-40.0999984741211}, {"数值"=timestamp(3724490076.000003 s since 1904-01-01), "数值 2"=-40.9000015258789}, {"数值"=timestamp(3724490176.000003 s since 1904-01-01), "数值 2"=-41.0}, {"数值"=timestamp(3724490276.000003 s since 1904-01-01), "数值 2"=-39.9000015258789}, {"数值"=timestamp(3724490376.000003 s since 1904-01-01), "数值 2"=-38.7000007629395}, {"数值"=timestamp(3724490476.000003 s since 1904-01-01), "数值 2"=-39.2000007629395}, {"数值"=timestamp(3724490576.000003 s since 1904-01-01), "数值 2"=-40.0999984741211}, {"数值"=timestamp(3724490676.000003 s since 1904-01-01), "数值 2"=-40.5999984741211}, {"数值"=timestamp(3724490776.000003 s since 1904-01-01), "数值 2"=-40.5999984741211}, {"数值"=timestamp(3724490876.000003 s since 1904-01-01), "数值 2"=-40.2000007629395}, {"数值"=timestamp(3724490976.000003 s since 1904-01-01), "数值 2"=-38.9000015258789}, {"数值"=timestamp(3724491076.000003 s since 1904-01-01), "数值 2"=-39.4000015258789}, {"数值"=timestamp(3724491176.000003 s since 1904-01-01), "数值 2"=-40.4000015258789}, {"数值"=timestamp(3724491276.000003 s since 1904-01-01), "数值 2"=-40.7000007629395}, {"数值"=timestamp(3724491376.000003 s since 1904-01-01), "数值 2"=-40.7000007629395}, {"数值"=timestamp(3724491476.000003 s since 1904-01-01), "数值 2"=62.7999992370605}, {"数值"=timestamp(3724491576.000003 s since 1904-01-01), "数值 2"=86.3000030517578}, {"数值"=timestamp(3724491676.000003 s since 1904-01-01), "数值 2"=85.1999969482422}, {"数值"=timestamp(3724491776.000003 s since 1904-01-01), "数值 2"=85.0999984741211}, {"数值"=timestamp(3724491876.000003 s since 1904-01-01), "数值 2"=85.0999984741211}, {"数值"=timestamp(3724491976.000003 s since 1904-01-01), "数值 2"=85.0}, {"数值"=timestamp(3724492076.000003 s since 1904-01-01), "数值 2"=85.0999984741211}, {"数值"=timestamp(3724492176.000003 s since 1904-01-01), "数值 2"=85.0}, {"数值"=timestamp(3724492276.000003 s since 1904-01-01), "数值 2"=85.0}, {"数值"=timestamp(3724492376.000003 s since 1904-01-01), "数值 2"=85.0}, {"数值"=timestamp(3724492476.000003 s since 1904-01-01), "数值 2"=85.0}, {"数值"=timestamp(3724492576.000003 s since 1904-01-01), "数值 2"=84.9000015258789}, {"数值"=timestamp(3724492676.000003 s since 1904-01-01), "数值 2"=85.0}, {"数值"=timestamp(3724492776.000003 s since 1904-01-01), "数值 2"=84.9000015258789}, {"数值"=timestamp(3724492876.000003 s since 1904-01-01), "数值 2"=84.9000015258789}, {"数值"=timestamp(3724492976.000003 s since 1904-01-01), "数值 2"=85.0}, {"数值"=timestamp(3724493076.000003 s since 1904-01-01), "数值 2"=84.9000015258789}, {"数值"=timestamp(3724493176.000003 s since 1904-01-01), "数值 2"=85.0999984741211}, {"数值"=timestamp(3724493276.000003 s since 1904-01-01), "数值 2"=-7.90000009536743}, {"数值"=timestamp(3724493376.000003 s since 1904-01-01), "数值 2"=-43.7000007629395}, {"数值"=timestamp(3724493476.000003 s since 1904-01-01), "数值 2"=-41.0}, {"数值"=timestamp(3724493576.000003 s since 1904-01-01), "数值 2"=-40.2999992370605}, {"数值"=timestamp(3724493676.000003 s since 1904-01-01), "数值 2"=-38.0}, {"数值"=timestamp(3724493776.000003 s since 1904-01-01), "数值 2"=-38.5999984741211}, {"数值"=timestamp(3724493876.000003 s since 1904-01-01), "数值 2"=-39.5}, {"数值"=timestamp(3724493976.000003 s since 1904-01-01), "数值 2"=-40.7999992370605}, {"数值"=timestamp(3724494076.000003 s since 1904-01-01), "数值 2"=-41.2000007629395}, {"数值"=timestamp(3724494176.000003 s since 1904-01-01), "数值 2"=-40.4000015258789}, {"数值"=timestamp(3724494276.000003 s since 1904-01-01), "数值 2"=-39.0}, {"数值"=timestamp(3724494376.000003 s since 1904-01-01), "数值 2"=-39.2999992370605}, {"数值"=timestamp(3724494476.000003 s since 1904-01-01), "数值 2"=-40.5}, {"数值"=timestamp(3724494576.000003 s since 1904-01-01), "数值 2"=-41.0999984741211}, {"数值"=timestamp(3724494676.000003 s since 1904-01-01), "数值 2"=-40.5}, {"数值"=timestamp(3724494776.000003 s since 1904-01-01), "数值 2"=-39.2000007629395}, {"数值"=timestamp(3724494876.000003 s since 1904-01-01), "数值 2"=-38.7000007629395}, {"数值"=timestamp(3724494976.000003 s since 1904-01-01), "数值 2"=-40.4000015258789}, {"数值"=timestamp(3724495076.000003 s since 1904-01-01), "数值 2"=-40.9000015258789}, {"数值"=timestamp(3724495176.000003 s since 1904-01-01), "数值 2"=-40.9000015258789}, {"数值"=timestamp(3724495276.000003 s since 1904-01-01), "数值 2"=-39.2000007629395}, {"数值"=timestamp(3724495376.000003 s since 1904-01-01), "数值 2"=-38.7000007629395}, {"数值"=timestamp(3724495476.000003 s since 1904-01-01), "数值 2"=-39.7000007629395}, {"数值"=timestamp(3724495576.000003 s since 1904-01-01), "数值 2"=-40.9000015258789}, {"数值"=timestamp(3724495676.000003 s since 1904-01-01), "数值 2"=-41.0999984741211}, {"数值"=timestamp(3724495776.000003 s since 1904-01-01), "数值 2"=-40.0999984741211}, {"数值"=timestamp(3724495876.000003 s since 1904-01-01), "数值 2"=-38.7000007629395}, {"数值"=timestamp(3724495976.000003 s since 1904-01-01), "数值 2"=78.1999969482422}, {"数值"=timestamp(3724496076.000003 s since 1904-01-01), "数值 2"=86.3000030517578}, {"数值"=timestamp(3724496176.000003 s since 1904-01-01), "数值 2"=85.0999984741211}, {"数值"=timestamp(3724496276.000003 s since 1904-01-01), "数值 2"=85.0}, {"数值"=timestamp(3724496376.000003 s since 1904-01-01), "数值 2"=85.0999984741211}, {"数值"=timestamp(3724496476.000003 s since 1904-01-01), "数值 2"=85.0}, {"数值"=timestamp(3724496576.000003 s since 1904-01-01), "数值 2"=85.0}, {"数值"=timestamp(3724496676.000003 s since 1904-01-01), "数值 2"=85.0}, {"数值"=timestamp(3724496776.000003 s since 1904-01-01), "数值 2"=85.0}, {"数值"=timestamp(3724496876.000003 s since 1904-01-01), "数值 2"=85.0999984741211}, {"数值"=timestamp(3724496976.000003 s since 1904-01-01), "数值 2"=84.9000015258789}, {"数值"=timestamp(3724497076.000003 s since 1904-01-01), "数值 2"=85.0999984741211}, {"数值"=timestamp(3724497176.000003 s since 1904-01-01), "数值 2"=85.0}, {"数值"=timestamp(3724497276.000003 s since 1904-01-01), "数值 2"=85.0999984741211}, {"数值"=timestamp(3724497376.000003 s since 1904-01-01), "数值 2"=85.0999984741211}, {"数值"=timestamp(3724497476.000003 s since 1904-01-01), "数值 2"=84.9000015258789}, {"数值"=timestamp(3724497576.000003 s since 1904-01-01), "数值 2"=85.0}, {"数值"=timestamp(3724497676.000003 s since 1904-01-01), "数值 2"=85.0999984741211}, {"数值"=timestamp(3724497776.000003 s since 1904-01-01), "数值 2"=-18.7000007629395}, {"数值"=timestamp(3724497876.000003 s since 1904-01-01), "数值 2"=-42.4000015258789}, {"数值"=timestamp(3724497976.000003 s since 1904-01-01), "数值 2"=-40.7000007629395}, {"数值"=timestamp(3724498076.000003 s since 1904-01-01), "数值 2"=-40.2000007629395}, {"数值"=timestamp(3724498176.000003 s since 1904-01-01), "数值 2"=-38.0}, {"数值"=timestamp(3724498276.000003 s since 1904-01-01), "数值 2"=-38.4000015258789}, {"数值"=timestamp(3724498376.000003 s since 1904-01-01), "数值 2"=-39.4000015258789}, {"数值"=timestamp(3724498476.000003 s since 1904-01-01), "数值 2"=-40.7000007629395}, {"数值"=timestamp(3724498576.000003 s since 1904-01-01), "数值 2"=-41.2000007629395}, {"数值"=timestamp(3724498676.000003 s since 1904-01-01), "数值 2"=-40.5999984741211}, {"数值"=timestamp(3724498776.000003 s since 1904-01-01), "数值 2"=-39.2999992370605}, {"数值"=timestamp(3724498876.000003 s since 1904-01-01), "数值 2"=-38.7000007629395}, {"数值"=timestamp(3724498976.000003 s since 1904-01-01), "数值 2"=-40.0}, {"数值"=timestamp(3724499076.000003 s since 1904-01-01), "数值 2"=-41.0}, {"数值"=timestamp(3724499176.000003 s since 1904-01-01), "数值 2"=-41.2000007629395}, {"数值"=timestamp(3724499276.000003 s since 1904-01-01), "数值 2"=-40.0999984741211}, {"数值"=timestamp(3724499376.000003 s since 1904-01-01), "数值 2"=-38.5999984741211}, {"数值"=timestamp(3724499476.000003 s since 1904-01-01), "数值 2"=-38.7999992370605}, {"数值"=timestamp(3724499576.000003 s since 1904-01-01), "数值 2"=-40.5999984741211}, {"数值"=timestamp(3724499676.000003 s since 1904-01-01), "数值 2"=-41.2000007629395}, {"数值"=timestamp(3724499776.000003 s since 1904-01-01), "数值 2"=-40.7999992370605}, {"数值"=timestamp(3724499876.000003 s since 1904-01-01), "数值 2"=-39.0999984741211}, {"数值"=timestamp(3724499976.000003 s since 1904-01-01), "数值 2"=-38.5999984741211}, {"数值"=timestamp(3724500076.000003 s since 1904-01-01), "数值 2"=-39.9000015258789}, {"数值"=timestamp(3724500176.000003 s since 1904-01-01), "数值 2"=-41.2000007629395}, {"数值"=timestamp(3724500276.000003 s since 1904-01-01), "数值 2"=-41.0}, {"数值"=timestamp(3724500376.000003 s since 1904-01-01), "数值 2"=-40.0999984741211}, {"数值"=timestamp(3724500476.000003 s since 1904-01-01), "数值 2"=86.6999969482422}, {"数值"=timestamp(3724500576.000003 s since 1904-01-01), "数值 2"=85.9000015258789}, {"数值"=timestamp(3724500676.000003 s since 1904-01-01), "数值 2"=85.0999984741211}, {"数值"=timestamp(3724500776.000003 s since 1904-01-01), "数值 2"=85.0999984741211}, {"数值"=timestamp(3724500876.000003 s since 1904-01-01), "数值 2"=85.0999984741211}, {"数值"=timestamp(3724500976.000003 s since 1904-01-01), "数值 2"=85.0}, {"数值"=timestamp(3724501076.000003 s since 1904-01-01), "数值 2"=85.0}, {"数值"=timestamp(3724501176.000003 s since 1904-01-01), "数值 2"=85.0}, {"数值"=timestamp(3724501276.000003 s since 1904-01-01), "数值 2"=85.0999984741211}, {"数值"=timestamp(3724501376.000003 s since 1904-01-01), "数值 2"=85.0999984741211}, {"数值"=timestamp(3724501476.000003 s since 1904-01-01), "数值 2"=85.0}, {"数值"=timestamp(3724501576.000003 s since 1904-01-01), "数值 2"=84.9000015258789}, {"数值"=timestamp(3724501676.000003 s since 1904-01-01), "数值 2"=85.0}, {"数值"=timestamp(3724501776.000003 s since 1904-01-01), "数值 2"=84.9000015258789}, {"数值"=timestamp(3724501876.000003 s since 1904-01-01), "数值 2"=84.9000015258789}, {"数值"=timestamp(3724501976.000003 s since 1904-01-01), "数值 2"=85.0999984741211}, {"数值"=timestamp(3724502076.000003 s since 1904-01-01), "数值 2"=85.0999984741211}, {"数值"=timestamp(3724502176.000003 s since 1904-01-01), "数值 2"=84.9000015258789}, {"数值"=timestamp(3724502276.000003 s since 1904-01-01), "数值 2"=-27.7999992370605}, {"数值"=timestamp(3724502376.000003 s since 1904-01-01), "数值 2"=-42.5999984741211}, {"数值"=timestamp(3724502476.000003 s since 1904-01-01), "数值 2"=-41.0999984741211}, {"数值"=timestamp(3724502576.000003 s since 1904-01-01), "数值 2"=-39.7999992370605}, {"数值"=timestamp(3724502676.000003 s since 1904-01-01), "数值 2"=-38.2000007629395}, {"数值"=timestamp(3724502776.000003 s since 1904-01-01), "数值 2"=-38.5}, {"数值"=timestamp(3724502876.000003 s since 1904-01-01), "数值 2"=-39.2000007629395}, {"数值"=timestamp(3724502976.000003 s since 1904-01-01), "数值 2"=-40.7999992370605}, {"数值"=timestamp(3724503076.000003 s since 1904-01-01), "数值 2"=-41.0999984741211}, {"数值"=timestamp(3724503176.000003 s since 1904-01-01), "数值 2"=-40.7999992370605}, {"数值"=timestamp(3724503276.000003 s since 1904-01-01), "数值 2"=-39.0999984741211}, {"数值"=timestamp(3724503376.000003 s since 1904-01-01), "数值 2"=-38.7000007629395}, {"数值"=timestamp(3724503476.000003 s since 1904-01-01), "数值 2"=-39.5999984741211}, {"数值"=timestamp(3724503576.000003 s since 1904-01-01), "数值 2"=-41.0}, {"数值"=timestamp(3724503676.000003 s since 1904-01-01), "数值 2"=-41.0999984741211}, {"数值"=timestamp(3724503776.000003 s since 1904-01-01), "数值 2"=-40.4000015258789}, {"数值"=timestamp(3724503876.000003 s since 1904-01-01), "数值 2"=-38.7000007629395}, {"数值"=timestamp(3724503976.000003 s since 1904-01-01), "数值 2"=-39.0}, {"数值"=timestamp(3724504076.000003 s since 1904-01-01), "数值 2"=-40.4000015258789}, {"数值"=timestamp(3724504176.000003 s since 1904-01-01), "数值 2"=-41.0999984741211}, {"数值"=timestamp(3724504276.000003 s since 1904-01-01), "数值 2"=-40.7000007629395}, {"数值"=timestamp(3724504376.000003 s since 1904-01-01), "数值 2"=-39.5999984741211}, {"数值"=timestamp(3724504476.000003 s since 1904-01-01), "数值 2"=-38.7000007629395}, {"数值"=timestamp(3724504576.000003 s since 1904-01-01), "数值 2"=-39.7000007629395}, {"数值"=timestamp(3724504676.000003 s since 1904-01-01), "数值 2"=-40.7999992370605}, {"数值"=timestamp(3724504776.000003 s since 1904-01-01), "数值 2"=-41.0}, {"数值"=timestamp(3724504876.000003 s since 1904-01-01), "数值 2"=-40.2999992370605}, {"数值"=timestamp(3724504976.000003 s since 1904-01-01), "数值 2"=36.2999992370605}, {"数值"=timestamp(3724505076.000003 s since 1904-01-01), "数值 2"=85.5}, {"数值"=timestamp(3724505176.000003 s since 1904-01-01), "数值 2"=85.0999984741211}, {"数值"=timestamp(3724505276.000003 s since 1904-01-01), "数值 2"=85.0}, {"数值"=timestamp(3724505376.000003 s since 1904-01-01), "数值 2"=85.0}, {"数值"=timestamp(3724505476.000003 s since 1904-01-01), "数值 2"=85.0}, {"数值"=timestamp(3724505576.000003 s since 1904-01-01), "数值 2"=85.0}, {"数值"=timestamp(3724505676.000003 s since 1904-01-01), "数值 2"=85.0999984741211}, {"数值"=timestamp(3724505776.000003 s since 1904-01-01), "数值 2"=85.0}, {"数值"=timestamp(3724505876.000003 s since 1904-01-01), "数值 2"=85.0}, {"数值"=timestamp(3724505976.000003 s since 1904-01-01), "数值 2"=85.0}, {"数值"=timestamp(3724506076.000003 s since 1904-01-01), "数值 2"=85.0}, {"数值"=timestamp(3724506176.000003 s since 1904-01-01), "数值 2"=85.0}, {"数值"=timestamp(3724506276.000003 s since 1904-01-01), "数值 2"=85.0}, {"数值"=timestamp(3724506376.000003 s since 1904-01-01), "数值 2"=85.0}, {"数值"=timestamp(3724506476.000003 s since 1904-01-01), "数值 2"=85.0999984741211}, {"数值"=timestamp(3724506576.000003 s since 1904-01-01), "数值 2"=84.9000015258789}, {"数值"=timestamp(3724506676.000003 s since 1904-01-01), "数值 2"=85.0}, {"数值"=timestamp(3724506776.000003 s since 1904-01-01), "数值 2"=13.3999996185303}, {"数值"=timestamp(3724506876.000003 s since 1904-01-01), "数值 2"=-41.5}, {"数值"=timestamp(3724506976.000003 s since 1904-01-01), "数值 2"=-40.5999984741211}, {"数值"=timestamp(3724507076.000003 s since 1904-01-01), "数值 2"=-40.2999992370605}, {"数值"=timestamp(3724507176.000003 s since 1904-01-01), "数值 2"=-38.0}, {"数值"=timestamp(3724507276.000003 s since 1904-01-01), "数值 2"=-38.5}, {"数值"=timestamp(3724507376.000003 s since 1904-01-01), "数值 2"=-39.2999992370605}, {"数值"=timestamp(3724507476.000003 s since 1904-01-01), "数值 2"=-40.5}, {"数值"=timestamp(3724507576.000003 s since 1904-01-01), "数值 2"=-41.0999984741211}, {"数值"=timestamp(3724507676.000003 s since 1904-01-01), "数值 2"=-40.7999992370605}, {"数值"=timestamp(3724507776.000003 s since 1904-01-01), "数值 2"=-39.4000015258789}, {"数值"=timestamp(3724507876.000003 s since 1904-01-01), "数值 2"=-38.5999984741211}, {"数值"=timestamp(3724507976.000003 s since 1904-01-01), "数值 2"=-39.5}, {"数值"=timestamp(3724508076.000003 s since 1904-01-01), "数值 2"=-40.9000015258789}, {"数值"=timestamp(3724508176.000003 s since 1904-01-01), "数值 2"=-41.0999984741211}, {"数值"=timestamp(3724508276.000003 s since 1904-01-01), "数值 2"=-40.5}, {"数值"=timestamp(3724508376.000003 s since 1904-01-01), "数值 2"=-38.7000007629395}, {"数值"=timestamp(3724508476.000003 s since 1904-01-01), "数值 2"=-38.9000015258789}, {"数值"=timestamp(3724508576.000003 s since 1904-01-01), "数值 2"=-40.2000007629395}, {"数值"=timestamp(3724508676.000003 s since 1904-01-01), "数值 2"=-41.0999984741211}, {"数值"=timestamp(3724508776.000003 s since 1904-01-01), "数值 2"=-40.9000015258789}, {"数值"=timestamp(3724508876.000003 s since 1904-01-01), "数值 2"=-39.7999992370605}, {"数值"=timestamp(3724508976.000003 s since 1904-01-01), "数值 2"=-38.5999984741211}, {"数值"=timestamp(3724509076.000003 s since 1904-01-01), "数值 2"=-39.2999992370605}, {"数值"=timestamp(3724509176.000003 s since 1904-01-01), "数值 2"=-40.7000007629395}, {"数值"=timestamp(3724509276.000003 s since 1904-01-01), "数值 2"=-41.2000007629395}, {"数值"=timestamp(3724509376.000003 s since 1904-01-01), "数值 2"=-40.5}, {"数值"=timestamp(3724509476.000003 s since 1904-01-01), "数值 2"=59.4000015258789}, {"数值"=timestamp(3724509576.000003 s since 1904-01-01), "数值 2"=85.1999969482422}, {"数值"=timestamp(3724509676.000003 s since 1904-01-01), "数值 2"=85.0}, {"数值"=timestamp(3724509776.000003 s since 1904-01-01), "数值 2"=85.0}, {"数值"=timestamp(3724509876.000003 s since 1904-01-01), "数值 2"=85.0}, {"数值"=timestamp(3724509976.000003 s since 1904-01-01), "数值 2"=85.0}, {"数值"=timestamp(3724510076.000003 s since 1904-01-01), "数值 2"=85.0}, {"数值"=timestamp(3724510176.000003 s since 1904-01-01), "数值 2"=85.0}, {"数值"=timestamp(3724510276.000003 s since 1904-01-01), "数值 2"=85.0}, {"数值"=timestamp(3724510376.000003 s since 1904-01-01), "数值 2"=85.0}, {"数值"=timestamp(3724510476.000003 s since 1904-01-01), "数值 2"=85.0}, {"数值"=timestamp(3724510576.000003 s since 1904-01-01), "数值 2"=84.9000015258789}, {"数值"=timestamp(3724510676.000003 s since 1904-01-01), "数值 2"=85.0}, {"数值"=timestamp(3724510776.000003 s since 1904-01-01), "数值 2"=85.0}, {"数值"=timestamp(3724510876.000003 s since 1904-01-01), "数值 2"=85.0}, {"数值"=timestamp(3724510976.000003 s since 1904-01-01), "数值 2"=85.0}, {"数值"=timestamp(3724511076.000003 s since 1904-01-01), "数值 2"=84.9000015258789}, {"数值"=timestamp(3724511176.000003 s since 1904-01-01), "数值 2"=85.0999984741211}, {"数值"=timestamp(3724511276.000003 s since 1904-01-01), "数值 2"=-4.40000009536743}, {"数值"=timestamp(3724511376.000003 s since 1904-01-01), "数值 2"=-43.2000007629395}, {"数值"=timestamp(3724511476.000003 s since 1904-01-01), "数值 2"=-40.9000015258789}, {"数值"=timestamp(3724511576.000003 s since 1904-01-01), "数值 2"=-40.0999984741211}, {"数值"=timestamp(3724511676.000003 s since 1904-01-01), "数值 2"=-38.0999984741211}, {"数值"=timestamp(3724511776.000003 s since 1904-01-01), "数值 2"=-38.7000007629395}, {"数值"=timestamp(3724511876.000003 s since 1904-01-01), "数值 2"=-39.5999984741211}, {"数值"=timestamp(3724511976.000003 s since 1904-01-01), "数值 2"=-40.7000007629395}, {"数值"=timestamp(3724512076.000003 s since 1904-01-01), "数值 2"=-41.0999984741211}, {"数值"=timestamp(3724512176.000003 s since 1904-01-01), "数值 2"=-40.5}, {"数值"=timestamp(3724512276.000003 s since 1904-01-01), "数值 2"=-39.0}, {"数值"=timestamp(3724512376.000003 s since 1904-01-01), "数值 2"=-39.0}, {"数值"=timestamp(3724512476.000003 s since 1904-01-01), "数值 2"=-40.5}, {"数值"=timestamp(3724512576.000003 s since 1904-01-01), "数值 2"=-41.0}, {"数值"=timestamp(3724512676.000003 s since 1904-01-01), "数值 2"=-40.7000007629395}, {"数值"=timestamp(3724512776.000003 s since 1904-01-01), "数值 2"=-39.4000015258789}, {"数值"=timestamp(3724512876.000003 s since 1904-01-01), "数值 2"=-38.5999984741211}, {"数值"=timestamp(3724512976.000003 s since 1904-01-01), "数值 2"=-40.0}, {"数值"=timestamp(3724513076.000003 s since 1904-01-01), "数值 2"=-40.9000015258789}, {"数值"=timestamp(3724513176.000003 s since 1904-01-01), "数值 2"=-41.0999984741211}, {"数值"=timestamp(3724513276.000003 s since 1904-01-01), "数值 2"=-40.0999984741211}, {"数值"=timestamp(3724513376.000003 s since 1904-01-01), "数值 2"=-38.7000007629395}, {"数值"=timestamp(3724513476.000003 s since 1904-01-01), "数值 2"=-38.9000015258789}, {"数值"=timestamp(3724513576.000003 s since 1904-01-01), "数值 2"=-40.5}, {"数值"=timestamp(3724513676.000003 s since 1904-01-01), "数值 2"=-41.0999984741211}, {"数值"=timestamp(3724513776.000003 s since 1904-01-01), "数值 2"=-40.9000015258789}, {"数值"=timestamp(3724513876.000003 s since 1904-01-01), "数值 2"=-39.4000015258789}, {"数值"=timestamp(3724513976.000003 s since 1904-01-01), "数值 2"=75.0999984741211}, {"数值"=timestamp(3724514076.000003 s since 1904-01-01), "数值 2"=86.4000015258789}, {"数值"=timestamp(3724514176.000003 s since 1904-01-01), "数值 2"=85.0}, {"数值"=timestamp(3724514276.000003 s since 1904-01-01), "数值 2"=85.0}, {"数值"=timestamp(3724514376.000003 s since 1904-01-01), "数值 2"=85.0999984741211}, {"数值"=timestamp(3724514476.000003 s since 1904-01-01), "数值 2"=85.0}, {"数值"=timestamp(3724514576.000003 s since 1904-01-01), "数值 2"=85.0}, {"数值"=timestamp(3724514676.000003 s since 1904-01-01), "数值 2"=85.0}, {"数值"=timestamp(3724514776.000003 s since 1904-01-01), "数值 2"=84.9000015258789}, {"数值"=timestamp(3724514876.000003 s since 1904-01-01), "数值 2"=84.9000015258789}, {"数值"=timestamp(3724514976.000003 s since 1904-01-01), "数值 2"=84.9000015258789}, {"数值"=timestamp(3724515076.000003 s since 1904-01-01), "数值 2"=85.0}, {"数值"=timestamp(3724515176.000003 s since 1904-01-01), "数值 2"=84.9000015258789}, {"数值"=timestamp(3724515276.000003 s since 1904-01-01), "数值 2"=84.9000015258789}, {"数值"=timestamp(3724515376.000003 s since 1904-01-01), "数值 2"=84.9000015258789}, {"数值"=timestamp(3724515476.000003 s since 1904-01-01), "数值 2"=85.0}, {"数值"=timestamp(3724515576.000003 s since 1904-01-01), "数值 2"=85.0}, {"数值"=timestamp(3724515676.000003 s since 1904-01-01), "数值 2"=84.9000015258789}, {"数值"=timestamp(3724515776.000003 s since 1904-01-01), "数值 2"=-16.1000003814697}, {"数值"=timestamp(3724515876.000003 s since 1904-01-01), "数值 2"=-42.7999992370605}, {"数值"=timestamp(3724515976.000003 s since 1904-01-01), "数值 2"=-40.7000007629395}, {"数值"=timestamp(3724516076.000003 s since 1904-01-01), "数值 2"=-40.0}, {"数值"=timestamp(3724516176.000003 s since 1904-01-01), "数值 2"=-38.0}, {"数值"=timestamp(3724516276.000003 s since 1904-01-01), "数值 2"=-38.9000015258789}, {"数值"=timestamp(3724516376.000003 s since 1904-01-01), "数值 2"=-39.7000007629395}, {"数值"=timestamp(3724516476.000003 s since 1904-01-01), "数值 2"=-40.7999992370605}, {"数值"=timestamp(3724516576.000003 s since 1904-01-01), "数值 2"=-41.0999984741211}, {"数值"=timestamp(3724516676.000003 s since 1904-01-01), "数值 2"=-40.4000015258789}, {"数值"=timestamp(3724516776.000003 s since 1904-01-01), "数值 2"=-39.0}, {"数值"=timestamp(3724516876.000003 s since 1904-01-01), "数值 2"=-38.7000007629395}, {"数值"=timestamp(3724516976.000003 s since 1904-01-01), "数值 2"=-40.5}, {"数值"=timestamp(3724517076.000003 s since 1904-01-01), "数值 2"=-41.0}, {"数值"=timestamp(3724517176.000003 s since 1904-01-01), "数值 2"=-40.9000015258789}, {"数值"=timestamp(3724517276.000003 s since 1904-01-01), "数值 2"=-39.5}, {"数值"=timestamp(3724517376.000003 s since 1904-01-01), "数值 2"=-38.7000007629395}, {"数值"=timestamp(3724517476.000003 s since 1904-01-01), "数值 2"=-39.5}, {"数值"=timestamp(3724517576.000003 s since 1904-01-01), "数值 2"=-41.0}, {"数值"=timestamp(3724517676.000003 s since 1904-01-01), "数值 2"=-41.0999984741211}, {"数值"=timestamp(3724517776.000003 s since 1904-01-01), "数值 2"=-40.2999992370605}, {"数值"=timestamp(3724517876.000003 s since 1904-01-01), "数值 2"=-38.5999984741211}, {"数值"=timestamp(3724517976.000003 s since 1904-01-01), "数值 2"=-38.9000015258789}, {"数值"=timestamp(3724518076.000003 s since 1904-01-01), "数值 2"=-40.5}, {"数值"=timestamp(3724518176.000003 s since 1904-01-01), "数值 2"=-41.2000007629395}, {"数值"=timestamp(3724518276.000003 s since 1904-01-01), "数值 2"=-40.7000007629395}, {"数值"=timestamp(3724518376.000003 s since 1904-01-01), "数值 2"=-39.2999992370605}, {"数值"=timestamp(3724518476.000003 s since 1904-01-01), "数值 2"=86.5}, {"数值"=timestamp(3724518576.000003 s since 1904-01-01), "数值 2"=85.9000015258789}, {"数值"=timestamp(3724518676.000003 s since 1904-01-01), "数值 2"=85.0999984741211}, {"数值"=timestamp(3724518776.000003 s since 1904-01-01), "数值 2"=85.0}, {"数值"=timestamp(3724518876.000003 s since 1904-01-01), "数值 2"=84.9000015258789}, {"数值"=timestamp(3724518976.000003 s since 1904-01-01), "数值 2"=85.0}, {"数值"=timestamp(3724519076.000003 s since 1904-01-01), "数值 2"=85.0}, {"数值"=timestamp(3724519176.000003 s since 1904-01-01), "数值 2"=85.0}, {"数值"=timestamp(3724519276.000003 s since 1904-01-01), "数值 2"=85.0999984741211}, {"数值"=timestamp(3724519376.000003 s since 1904-01-01), "数值 2"=84.9000015258789}, {"数值"=timestamp(3724519476.000003 s since 1904-01-01), "数值 2"=85.0}, {"数值"=timestamp(3724519576.000003 s since 1904-01-01), "数值 2"=85.0}, {"数值"=timestamp(3724519676.000003 s since 1904-01-01), "数值 2"=85.0}, {"数值"=timestamp(3724519776.000003 s since 1904-01-01), "数值 2"=85.0999984741211}, {"数值"=timestamp(3724519876.000003 s since 1904-01-01), "数值 2"=85.0}, {"数值"=timestamp(3724519976.000003 s since 1904-01-01), "数值 2"=85.0}, {"数值"=timestamp(3724520076.000003 s since 1904-01-01), "数值 2"=85.0999984741211}, {"数值"=timestamp(3724520176.000003 s since 1904-01-01), "数值 2"=85.0}, {"数值"=timestamp(3724520276.000003 s since 1904-01-01), "数值 2"=-24.0}, {"数值"=timestamp(3724520376.000003 s since 1904-01-01), "数值 2"=-42.0}, {"数值"=timestamp(3724520476.000003 s since 1904-01-01), "数值 2"=-40.7000007629395}, {"数值"=timestamp(3724520576.000003 s since 1904-01-01), "数值 2"=-40.2000007629395}, {"数值"=timestamp(3724520676.000003 s since 1904-01-01), "数值 2"=-37.9000015258789}, {"数值"=timestamp(3724520776.000003 s since 1904-01-01), "数值 2"=-38.4000015258789}, {"数值"=timestamp(3724520876.000003 s since 1904-01-01), "数值 2"=-39.5999984741211}, {"数值"=timestamp(3724520976.000003 s since 1904-01-01), "数值 2"=-40.7000007629395}, {"数值"=timestamp(3724521076.000003 s since 1904-01-01), "数值 2"=-41.2000007629395}, {"数值"=timestamp(3724521176.000003 s since 1904-01-01), "数值 2"=-40.5999984741211}, {"数值"=timestamp(3724521276.000003 s since 1904-01-01), "数值 2"=-39.4000015258789}, {"数值"=timestamp(3724521376.000003 s since 1904-01-01), "数值 2"=-38.5999984741211}, {"数值"=timestamp(3724521476.000003 s since 1904-01-01), "数值 2"=-40.0999984741211}, {"数值"=timestamp(3724521576.000003 s since 1904-01-01), "数值 2"=-40.9000015258789}, {"数值"=timestamp(3724521676.000003 s since 1904-01-01), "数值 2"=-41.0999984741211}, {"数值"=timestamp(3724521776.000003 s since 1904-01-01), "数值 2"=-40.0999984741211}, {"数值"=timestamp(3724521876.000003 s since 1904-01-01), "数值 2"=-38.7000007629395}, {"数值"=timestamp(3724521976.000003 s since 1904-01-01), "数值 2"=-38.9000015258789}, {"数值"=timestamp(3724522076.000003 s since 1904-01-01), "数值 2"=-40.7000007629395}, {"数值"=timestamp(3724522176.000003 s since 1904-01-01), "数值 2"=-41.0999984741211}, {"数值"=timestamp(3724522276.000003 s since 1904-01-01), "数值 2"=-40.7000007629395}, {"数值"=timestamp(3724522376.000003 s since 1904-01-01), "数值 2"=-39.0999984741211}, {"数值"=timestamp(3724522476.000003 s since 1904-01-01), "数值 2"=-38.7000007629395}, {"数值"=timestamp(3724522576.000003 s since 1904-01-01), "数值 2"=-39.7000007629395}, {"数值"=timestamp(3724522676.000003 s since 1904-01-01), "数值 2"=-41.0}, {"数值"=timestamp(3724522776.000003 s since 1904-01-01), "数值 2"=-41.0}, {"数值"=timestamp(3724522876.000003 s since 1904-01-01), "数值 2"=-40.0999984741211}, {"数值"=timestamp(3724522976.000003 s since 1904-01-01), "数值 2"=90.3000030517578}, {"数值"=timestamp(3724523076.000003 s since 1904-01-01), "数值 2"=85.5999984741211}, {"数值"=timestamp(3724523176.000003 s since 1904-01-01), "数值 2"=85.0}, {"数值"=timestamp(3724523276.000003 s since 1904-01-01), "数值 2"=85.0}, {"数值"=timestamp(3724523376.000003 s since 1904-01-01), "数值 2"=85.0}, {"数值"=timestamp(3724523476.000003 s since 1904-01-01), "数值 2"=85.0}, {"数值"=timestamp(3724523576.000003 s since 1904-01-01), "数值 2"=85.0999984741211}, {"数值"=timestamp(3724523676.000003 s since 1904-01-01), "数值 2"=85.0999984741211}, {"数值"=timestamp(3724523776.000003 s since 1904-01-01), "数值 2"=84.9000015258789}, {"数值"=timestamp(3724523876.000003 s since 1904-01-01), "数值 2"=85.0999984741211}, {"数值"=timestamp(3724523976.000003 s since 1904-01-01), "数值 2"=85.0999984741211}, {"数值"=timestamp(3724524076.000003 s since 1904-01-01), "数值 2"=85.0}, {"数值"=timestamp(3724524176.000003 s since 1904-01-01), "数值 2"=85.0}, {"数值"=timestamp(3724524276.000003 s since 1904-01-01), "数值 2"=85.0}, {"数值"=timestamp(3724524376.000003 s since 1904-01-01), "数值 2"=85.0999984741211}, {"数值"=timestamp(3724524476.000003 s since 1904-01-01), "数值 2"=84.9000015258789}, {"数值"=timestamp(3724524576.000003 s since 1904-01-01), "数值 2"=85.0999984741211}, {"数值"=timestamp(3724524676.000003 s since 1904-01-01), "数值 2"=85.0}, {"数值"=timestamp(3724524776.000003 s since 1904-01-01), "数值 2"=19.2000007629395}, {"数值"=timestamp(3724524876.000003 s since 1904-01-01), "数值 2"=-42.2999992370605}, {"数值"=timestamp(3724524976.000003 s since 1904-01-01), "数值 2"=-40.7999992370605}, {"数值"=timestamp(3724525076.000003 s since 1904-01-01), "数值 2"=-40.5}, {"数值"=timestamp(3724525176.000003 s since 1904-01-01), "数值 2"=-38.0}, {"数值"=timestamp(3724525276.000003 s since 1904-01-01), "数值 2"=-38.4000015258789}, {"数值"=timestamp(3724525376.000003 s since 1904-01-01), "数值 2"=-39.2999992370605}, {"数值"=timestamp(3724525476.000003 s since 1904-01-01), "数值 2"=-40.9000015258789}, {"数值"=timestamp(3724525576.000003 s since 1904-01-01), "数值 2"=-41.0}, {"数值"=timestamp(3724525676.000003 s since 1904-01-01), "数值 2"=-40.5999984741211}, {"数值"=timestamp(3724525776.000003 s since 1904-01-01), "数值 2"=-38.9000015258789}, {"数值"=timestamp(3724525876.000003 s since 1904-01-01), "数值 2"=-38.7999992370605}, {"数值"=timestamp(3724525976.000003 s since 1904-01-01), "数值 2"=-40.4000015258789}, {"数值"=timestamp(3724526076.000003 s since 1904-01-01), "数值 2"=-41.0}, {"数值"=timestamp(3724526176.000003 s since 1904-01-01), "数值 2"=-40.7999992370605}, {"数值"=timestamp(3724526276.000003 s since 1904-01-01), "数值 2"=-39.5}, {"数值"=timestamp(3724526376.000003 s since 1904-01-01), "数值 2"=-38.7000007629395}, {"数值"=timestamp(3724526476.000003 s since 1904-01-01), "数值 2"=-40.0999984741211}, {"数值"=timestamp(3724526576.000003 s since 1904-01-01), "数值 2"=-40.7999992370605}, {"数值"=timestamp(3724526676.000003 s since 1904-01-01), "数值 2"=-40.9000015258789}, {"数值"=timestamp(3724526776.000003 s since 1904-01-01), "数值 2"=-40.0}, {"数值"=timestamp(3724526876.000003 s since 1904-01-01), "数值 2"=-38.7000007629395}, {"数值"=timestamp(3724526976.000003 s since 1904-01-01), "数值 2"=-39.5}, {"数值"=timestamp(3724527076.000003 s since 1904-01-01), "数值 2"=-40.7999992370605}, {"数值"=timestamp(3724527176.000003 s since 1904-01-01), "数值 2"=-41.0999984741211}, {"数值"=timestamp(3724527276.000003 s since 1904-01-01), "数值 2"=-40.4000015258789}, {"数值"=timestamp(3724527376.000003 s since 1904-01-01), "数值 2"=-39.0}, {"数值"=timestamp(3724527476.000003 s since 1904-01-01), "数值 2"=55.5999984741211}, {"数值"=timestamp(3724527576.000003 s since 1904-01-01), "数值 2"=85.3000030517578}, {"数值"=timestamp(3724527676.000003 s since 1904-01-01), "数值 2"=85.0}, {"数值"=timestamp(3724527776.000003 s since 1904-01-01), "数值 2"=85.0}, {"数值"=timestamp(3724527876.000003 s since 1904-01-01), "数值 2"=85.0}, {"数值"=timestamp(3724527976.000003 s since 1904-01-01), "数值 2"=85.0}, {"数值"=timestamp(3724528076.000003 s since 1904-01-01), "数值 2"=85.0}, {"数值"=timestamp(3724528176.000003 s since 1904-01-01), "数值 2"=85.0}, {"数值"=timestamp(3724528276.000003 s since 1904-01-01), "数值 2"=85.0999984741211}, {"数值"=timestamp(3724528376.000003 s since 1904-01-01), "数值 2"=84.9000015258789}, {"数值"=timestamp(3724528476.000003 s since 1904-01-01), "数值 2"=85.0}, {"数值"=timestamp(3724528576.000003 s since 1904-01-01), "数值 2"=85.0}, {"数值"=timestamp(3724528676.000003 s since 1904-01-01), "数值 2"=84.9000015258789}, {"数值"=timestamp(3724528776.000003 s since 1904-01-01), "数值 2"=85.0}, {"数值"=timestamp(3724528876.000003 s since 1904-01-01), "数值 2"=85.0999984741211}, {"数值"=timestamp(3724528976.000003 s since 1904-01-01), "数值 2"=85.0}, {"数值"=timestamp(3724529076.000003 s since 1904-01-01), "数值 2"=85.0}, {"数值"=timestamp(3724529176.000003 s since 1904-01-01), "数值 2"=85.0999984741211}, {"数值"=timestamp(3724529276.000003 s since 1904-01-01), "数值 2"=3.20000004768372}, {"数值"=timestamp(3724529376.000003 s since 1904-01-01), "数值 2"=-42.0}, {"数值"=timestamp(3724529476.000003 s since 1904-01-01), "数值 2"=-40.7000007629395}, {"数值"=timestamp(3724529576.000003 s since 1904-01-01), "数值 2"=-40.0999984741211}, {"数值"=timestamp(3724529676.000003 s since 1904-01-01), "数值 2"=-38.0}, {"数值"=timestamp(3724529776.000003 s since 1904-01-01), "数值 2"=-38.5999984741211}, {"数值"=timestamp(3724529876.000003 s since 1904-01-01), "数值 2"=-39.5}, {"数值"=timestamp(3724529976.000003 s since 1904-01-01), "数值 2"=-40.9000015258789}, {"数值"=timestamp(3724530076.000003 s since 1904-01-01), "数值 2"=-41.0999984741211}, {"数值"=timestamp(3724530176.000003 s since 1904-01-01), "数值 2"=-40.5}, {"数值"=timestamp(3724530276.000003 s since 1904-01-01), "数值 2"=-38.7000007629395}, {"数值"=timestamp(3724530376.000003 s since 1904-01-01), "数值 2"=-38.9000015258789}, {"数值"=timestamp(3724530476.000003 s since 1904-01-01), "数值 2"=-40.4000015258789}, {"数值"=timestamp(3724530576.000003 s since 1904-01-01), "数值 2"=-41.0}, {"数值"=timestamp(3724530676.000003 s since 1904-01-01), "数值 2"=-40.7999992370605}, {"数值"=timestamp(3724530776.000003 s since 1904-01-01), "数值 2"=-39.7000007629395}, {"数值"=timestamp(3724530876.000003 s since 1904-01-01), "数值 2"=-38.5999984741211}, {"数值"=timestamp(3724530976.000003 s since 1904-01-01), "数值 2"=-40.0}, {"数值"=timestamp(3724531076.000003 s since 1904-01-01), "数值 2"=-40.7999992370605}, {"数值"=timestamp(3724531176.000003 s since 1904-01-01), "数值 2"=-41.0}, {"数值"=timestamp(3724531276.000003 s since 1904-01-01), "数值 2"=-40.0}, {"数值"=timestamp(3724531376.000003 s since 1904-01-01), "数值 2"=-38.5999984741211}, {"数值"=timestamp(3724531476.000003 s since 1904-01-01), "数值 2"=-38.9000015258789}, {"数值"=timestamp(3724531576.000003 s since 1904-01-01), "数值 2"=-40.7000007629395}, {"数值"=timestamp(3724531676.000003 s since 1904-01-01), "数值 2"=-41.2000007629395}, {"数值"=timestamp(3724531776.000003 s since 1904-01-01), "数值 2"=-40.7000007629395}, {"数值"=timestamp(3724531876.000003 s since 1904-01-01), "数值 2"=-38.9000015258789}, {"数值"=timestamp(3724531976.000003 s since 1904-01-01), "数值 2"=71.9000015258789}, {"数值"=timestamp(3724532076.000003 s since 1904-01-01), "数值 2"=86.3000030517578}, {"数值"=timestamp(3724532176.000003 s since 1904-01-01), "数值 2"=85.0999984741211}, {"数值"=timestamp(3724532276.000003 s since 1904-01-01), "数值 2"=85.0}, {"数值"=timestamp(3724532376.000003 s since 1904-01-01), "数值 2"=85.0}, {"数值"=timestamp(3724532476.000003 s since 1904-01-01), "数值 2"=85.0}, {"数值"=timestamp(3724532576.000003 s since 1904-01-01), "数值 2"=85.0}, {"数值"=timestamp(3724532676.000003 s since 1904-01-01), "数值 2"=85.0}, {"数值"=timestamp(3724532776.000003 s since 1904-01-01), "数值 2"=85.0999984741211}, {"数值"=timestamp(3724532876.000003 s since 1904-01-01), "数值 2"=85.0}, {"数值"=timestamp(3724532976.000003 s since 1904-01-01), "数值 2"=85.0}, {"数值"=timestamp(3724533076.000003 s since 1904-01-01), "数值 2"=85.0}, {"数值"=timestamp(3724533176.000003 s since 1904-01-01), "数值 2"=85.0}, {"数值"=timestamp(3724533276.000003 s since 1904-01-01), "数值 2"=85.0}, {"数值"=timestamp(3724533376.000003 s since 1904-01-01), "数值 2"=85.0999984741211}, {"数值"=timestamp(3724533476.000003 s since 1904-01-01), "数值 2"=85.0}, {"数值"=timestamp(3724533576.000003 s since 1904-01-01), "数值 2"=84.9000015258789}, {"数值"=timestamp(3724533676.000003 s since 1904-01-01), "数值 2"=85.0}, {"数值"=timestamp(3724533776.000003 s since 1904-01-01), "数值 2"=-12.6000003814697}, {"数值"=timestamp(3724533876.000003 s since 1904-01-01), "数值 2"=-43.5}, {"数值"=timestamp(3724533976.000003 s since 1904-01-01), "数值 2"=-40.7999992370605}, {"数值"=timestamp(3724534076.000003 s since 1904-01-01), "数值 2"=-40.0}, {"数值"=timestamp(3724534176.000003 s since 1904-01-01), "数值 2"=-38.0999984741211}, {"数值"=timestamp(3724534276.000003 s since 1904-01-01), "数值 2"=-38.7999992370605}, {"数值"=timestamp(3724534376.000003 s since 1904-01-01), "数值 2"=-39.4000015258789}, {"数值"=timestamp(3724534476.000003 s since 1904-01-01), "数值 2"=-40.5999984741211}, {"数值"=timestamp(3724534576.000003 s since 1904-01-01), "数值 2"=-41.0999984741211}, {"数值"=timestamp(3724534676.000003 s since 1904-01-01), "数值 2"=-40.7000007629395}, {"数值"=timestamp(3724534776.000003 s since 1904-01-01), "数值 2"=-39.2999992370605}, {"数值"=timestamp(3724534876.000003 s since 1904-01-01), "数值 2"=-38.7999992370605}, {"数值"=timestamp(3724534976.000003 s since 1904-01-01), "数值 2"=-40.0}, {"数值"=timestamp(3724535076.000003 s since 1904-01-01), "数值 2"=-41.0}, {"数值"=timestamp(3724535176.000003 s since 1904-01-01), "数值 2"=-41.0}, {"数值"=timestamp(3724535276.000003 s since 1904-01-01), "数值 2"=-40.0}, {"数值"=timestamp(3724535376.000003 s since 1904-01-01), "数值 2"=-38.5999984741211}, {"数值"=timestamp(3724535476.000003 s since 1904-01-01), "数值 2"=-39.0999984741211}, {"数值"=timestamp(3724535576.000003 s since 1904-01-01), "数值 2"=-40.7000007629395}, {"数值"=timestamp(3724535676.000003 s since 1904-01-01), "数值 2"=-41.2000007629395}, {"数值"=timestamp(3724535776.000003 s since 1904-01-01), "数值 2"=-40.7000007629395}, {"数值"=timestamp(3724535876.000003 s since 1904-01-01), "数值 2"=-39.2999992370605}, {"数值"=timestamp(3724535976.000003 s since 1904-01-01), "数值 2"=-38.5999984741211}, {"数值"=timestamp(3724536076.000003 s since 1904-01-01), "数值 2"=-39.7999992370605}, {"数值"=timestamp(3724536176.000003 s since 1904-01-01), "数值 2"=-40.9000015258789}, {"数值"=timestamp(3724536276.000003 s since 1904-01-01), "数值 2"=-41.2999992370605}, {"数值"=timestamp(3724536376.000003 s since 1904-01-01), "数值 2"=-40.4000015258789}, {"数值"=timestamp(3724536476.000003 s since 1904-01-01), "数值 2"=81.4000015258789}, {"数值"=timestamp(3724536576.000003 s since 1904-01-01), "数值 2"=86.1999969482422}, {"数值"=timestamp(3724536676.000003 s since 1904-01-01), "数值 2"=85.1999969482422}, {"数值"=timestamp(3724536776.000003 s since 1904-01-01), "数值 2"=85.0}, {"数值"=timestamp(3724536876.000003 s since 1904-01-01), "数值 2"=85.0999984741211}, {"数值"=timestamp(3724536976.000003 s since 1904-01-01), "数值 2"=84.9000015258789}, {"数值"=timestamp(3724537076.000003 s since 1904-01-01), "数值 2"=85.0}, {"数值"=timestamp(3724537176.000003 s since 1904-01-01), "数值 2"=85.0}, {"数值"=timestamp(3724537276.000003 s since 1904-01-01), "数值 2"=85.0}, {"数值"=timestamp(3724537376.000003 s since 1904-01-01), "数值 2"=85.0999984741211}, {"数值"=timestamp(3724537476.000003 s since 1904-01-01), "数值 2"=85.0999984741211}, {"数值"=timestamp(3724537576.000003 s since 1904-01-01), "数值 2"=85.0}, {"数值"=timestamp(3724537676.000003 s since 1904-01-01), "数值 2"=85.0}, {"数值"=timestamp(3724537776.000003 s since 1904-01-01), "数值 2"=85.0999984741211}, {"数值"=timestamp(3724537876.000003 s since 1904-01-01), "数值 2"=85.0}, {"数值"=timestamp(3724537976.000003 s since 1904-01-01), "数值 2"=85.0}, {"数值"=timestamp(3724538076.000003 s since 1904-01-01), "数值 2"=85.0}, {"数值"=timestamp(3724538176.000003 s since 1904-01-01), "数值 2"=85.0999984741211}, {"数值"=timestamp(3724538276.000003 s since 1904-01-01), "数值 2"=-22.8999996185303}, {"数值"=timestamp(3724538376.000003 s since 1904-01-01), "数值 2"=-41.9000015258789}, {"数值"=timestamp(3724538476.000003 s since 1904-01-01), "数值 2"=-40.5999984741211}, {"数值"=timestamp(3724538576.000003 s since 1904-01-01), "数值 2"=-40.2000007629395}, {"数值"=timestamp(3724538676.000003 s since 1904-01-01), "数值 2"=-38.0}, {"数值"=timestamp(3724538776.000003 s since 1904-01-01), "数值 2"=-38.2999992370605}, {"数值"=timestamp(3724538876.000003 s since 1904-01-01), "数值 2"=-39.5}, {"数值"=timestamp(3724538976.000003 s since 1904-01-01), "数值 2"=-40.7000007629395}, {"数值"=timestamp(3724539076.000003 s since 1904-01-01), "数值 2"=-41.4000015258789}, {"数值"=timestamp(3724539176.000003 s since 1904-01-01), "数值 2"=-40.9000015258789}, {"数值"=timestamp(3724539276.000003 s since 1904-01-01), "数值 2"=-39.5999984741211}, {"数值"=timestamp(3724539376.000003 s since 1904-01-01), "数值 2"=-38.5}, {"数值"=timestamp(3724539476.000003 s since 1904-01-01), "数值 2"=-39.5999984741211}, {"数值"=timestamp(3724539576.000003 s since 1904-01-01), "数值 2"=-40.7999992370605}, {"数值"=timestamp(3724539676.000003 s since 1904-01-01), "数值 2"=-41.0999984741211}, {"数值"=timestamp(3724539776.000003 s since 1904-01-01), "数值 2"=-40.2000007629395}, {"数值"=timestamp(3724539876.000003 s since 1904-01-01), "数值 2"=-38.7000007629395}, {"数值"=timestamp(3724539976.000003 s since 1904-01-01), "数值 2"=-38.7000007629395}, {"数值"=timestamp(3724540076.000003 s since 1904-01-01), "数值 2"=-40.5999984741211}, {"数值"=timestamp(3724540176.000003 s since 1904-01-01), "数值 2"=-41.0999984741211}, {"数值"=timestamp(3724540276.000003 s since 1904-01-01), "数值 2"=-40.9000015258789}, {"数值"=timestamp(3724540376.000003 s since 1904-01-01), "数值 2"=-39.2000007629395}, {"数值"=timestamp(3724540476.000003 s since 1904-01-01), "数值 2"=-38.7000007629395}, {"数值"=timestamp(3724540576.000003 s since 1904-01-01), "数值 2"=-39.5999984741211}, {"数值"=timestamp(3724540676.000003 s since 1904-01-01), "数值 2"=-41.0}, {"数值"=timestamp(3724540776.000003 s since 1904-01-01), "数值 2"=-41.0999984741211}, {"数值"=timestamp(3724540876.000003 s since 1904-01-01), "数值 2"=-40.2000007629395}, {"数值"=timestamp(3724540976.000003 s since 1904-01-01), "数值 2"=87.5999984741211}, {"数值"=timestamp(3724541076.000003 s since 1904-01-01), "数值 2"=85.9000015258789}, {"数值"=timestamp(3724541176.000003 s since 1904-01-01), "数值 2"=85.3000030517578}, {"数值"=timestamp(3724541276.000003 s since 1904-01-01), "数值 2"=85.0999984741211}, {"数值"=timestamp(3724541376.000003 s since 1904-01-01), "数值 2"=84.9000015258789}, {"数值"=timestamp(3724541476.000003 s since 1904-01-01), "数值 2"=85.0}, {"数值"=timestamp(3724541576.000003 s since 1904-01-01), "数值 2"=85.0}, {"数值"=timestamp(3724541676.000003 s since 1904-01-01), "数值 2"=85.0}, {"数值"=timestamp(3724541776.000003 s since 1904-01-01), "数值 2"=85.0}, {"数值"=timestamp(3724541876.000003 s since 1904-01-01), "数值 2"=85.0999984741211}, {"数值"=timestamp(3724541976.000003 s since 1904-01-01), "数值 2"=85.0}, {"数值"=timestamp(3724542076.000003 s since 1904-01-01), "数值 2"=85.0}, {"数值"=timestamp(3724542176.000003 s since 1904-01-01), "数值 2"=85.0}, {"数值"=timestamp(3724542276.000003 s since 1904-01-01), "数值 2"=85.0}, {"数值"=timestamp(3724542376.000003 s since 1904-01-01), "数值 2"=85.0999984741211}, {"数值"=timestamp(3724542476.000003 s since 1904-01-01), "数值 2"=85.0}, {"数值"=timestamp(3724542576.000003 s since 1904-01-01), "数值 2"=84.9000015258789}, {"数值"=timestamp(3724542676.000003 s since 1904-01-01), "数值 2"=85.0999984741211}, {"数值"=timestamp(3724542776.000003 s since 1904-01-01), "数值 2"=-29.3999996185303}, {"数值"=timestamp(3724542876.000003 s since 1904-01-01), "数值 2"=-42.0}, {"数值"=timestamp(3724542976.000003 s since 1904-01-01), "数值 2"=-40.7000007629395}, {"数值"=timestamp(3724543076.000003 s since 1904-01-01), "数值 2"=-39.7999992370605}, {"数值"=timestamp(3724543176.000003 s since 1904-01-01), "数值 2"=-37.7999992370605}, {"数值"=timestamp(3724543276.000003 s since 1904-01-01), "数值 2"=-38.2999992370605}, {"数值"=timestamp(3724543376.000003 s since 1904-01-01), "数值 2"=-39.7000007629395}, {"数值"=timestamp(3724543476.000003 s since 1904-01-01), "数值 2"=-40.5}, {"数值"=timestamp(3724543576.000003 s since 1904-01-01), "数值 2"=-40.7999992370605}, {"数值"=timestamp(3724543676.000003 s since 1904-01-01), "数值 2"=-40.7000007629395}, {"数值"=timestamp(3724543776.000003 s since 1904-01-01), "数值 2"=-39.4000015258789}, {"数值"=timestamp(3724543876.000003 s since 1904-01-01), "数值 2"=-38.7999992370605}, {"数值"=timestamp(3724543976.000003 s since 1904-01-01), "数值 2"=-40.5}, {"数值"=timestamp(3724544076.000003 s since 1904-01-01), "数值 2"=-41.2000007629395}, {"数值"=timestamp(3724544176.000003 s since 1904-01-01), "数值 2"=-41.0999984741211}, {"数值"=timestamp(3724544276.000003 s since 1904-01-01), "数值 2"=-39.7000007629395}, {"数值"=timestamp(3724544376.000003 s since 1904-01-01), "数值 2"=-38.4000015258789}, {"数值"=timestamp(3724544476.000003 s since 1904-01-01), "数值 2"=-38.9000015258789}, {"数值"=timestamp(3724544576.000003 s since 1904-01-01), "数值 2"=-40.7999992370605}, {"数值"=timestamp(3724544676.000003 s since 1904-01-01), "数值 2"=-41.0999984741211}, {"数值"=timestamp(3724544776.000003 s since 1904-01-01), "数值 2"=-40.5999984741211}, {"数值"=timestamp(3724544876.000003 s since 1904-01-01), "数值 2"=-38.7000007629395}, {"数值"=timestamp(3724544976.000003 s since 1904-01-01), "数值 2"=-38.7999992370605}, {"数值"=timestamp(3724545076.000003 s since 1904-01-01), "数值 2"=-40.4000015258789}, {"数值"=timestamp(3724545176.000003 s since 1904-01-01), "数值 2"=-41.2000007629395}, {"数值"=timestamp(3724545276.000003 s since 1904-01-01), "数值 2"=-40.7000007629395}, {"数值"=timestamp(3724545376.000003 s since 1904-01-01), "数值 2"=-39.4000015258789}, {"数值"=timestamp(3724545476.000003 s since 1904-01-01), "数值 2"=50.7000007629395}, {"数值"=timestamp(3724545576.000003 s since 1904-01-01), "数值 2"=85.5999984741211}, {"数值"=timestamp(3724545676.000003 s since 1904-01-01), "数值 2"=85.1999969482422}, {"数值"=timestamp(3724545776.000003 s since 1904-01-01), "数值 2"=85.0999984741211}, {"数值"=timestamp(3724545876.000003 s since 1904-01-01), "数值 2"=85.0999984741211}, {"数值"=timestamp(3724545976.000003 s since 1904-01-01), "数值 2"=84.9000015258789}, {"数值"=timestamp(3724546076.000003 s since 1904-01-01), "数值 2"=85.0}, {"数值"=timestamp(3724546176.000003 s since 1904-01-01), "数值 2"=85.0}, {"数值"=timestamp(3724546276.000003 s since 1904-01-01), "数值 2"=85.0}, {"数值"=timestamp(3724546376.000003 s since 1904-01-01), "数值 2"=85.0}, {"数值"=timestamp(3724546476.000003 s since 1904-01-01), "数值 2"=85.0999984741211}, {"数值"=timestamp(3724546576.000003 s since 1904-01-01), "数值 2"=84.9000015258789}, {"数值"=timestamp(3724546676.000003 s since 1904-01-01), "数值 2"=85.0999984741211}, {"数值"=timestamp(3724546776.000003 s since 1904-01-01), "数值 2"=85.0}, {"数值"=timestamp(3724546876.000003 s since 1904-01-01), "数值 2"=85.0}, {"数值"=timestamp(3724546976.000003 s since 1904-01-01), "数值 2"=85.0999984741211}, {"数值"=timestamp(3724547076.000003 s since 1904-01-01), "数值 2"=84.9000015258789}, {"数值"=timestamp(3724547176.000003 s since 1904-01-01), "数值 2"=85.0}, {"数值"=timestamp(3724547276.000003 s since 1904-01-01), "数值 2"=2.40000009536743}, {"数值"=timestamp(3724547376.000003 s since 1904-01-01), "数值 2"=-42.2000007629395}, {"数值"=timestamp(3724547476.000003 s since 1904-01-01), "数值 2"=-41.0}, {"数值"=timestamp(3724547576.000003 s since 1904-01-01), "数值 2"=-40.2000007629395}, {"数值"=timestamp(3724547676.000003 s since 1904-01-01), "数值 2"=-38.0}, {"数值"=timestamp(3724547776.000003 s since 1904-01-01), "数值 2"=-38.5}, {"数值"=timestamp(3724547876.000003 s since 1904-01-01), "数值 2"=-39.7000007629395}, {"数值"=timestamp(3724547976.000003 s since 1904-01-01), "数值 2"=-40.7999992370605}, {"数值"=timestamp(3724548076.000003 s since 1904-01-01), "数值 2"=-40.7000007629395}, {"数值"=timestamp(3724548176.000003 s since 1904-01-01), "数值 2"=-40.5999984741211}, {"数值"=timestamp(3724548276.000003 s since 1904-01-01), "数值 2"=-38.9000015258789}, {"数值"=timestamp(3724548376.000003 s since 1904-01-01), "数值 2"=-38.9000015258789}, {"数值"=timestamp(3724548476.000003 s since 1904-01-01), "数值 2"=-40.4000015258789}, {"数值"=timestamp(3724548576.000003 s since 1904-01-01), "数值 2"=-41.0999984741211}, {"数值"=timestamp(3724548676.000003 s since 1904-01-01), "数值 2"=-40.7999992370605}, {"数值"=timestamp(3724548776.000003 s since 1904-01-01), "数值 2"=-39.5}, {"数值"=timestamp(3724548876.000003 s since 1904-01-01), "数值 2"=-38.7000007629395}, {"数值"=timestamp(3724548976.000003 s since 1904-01-01), "数值 2"=-40.2999992370605}, {"数值"=timestamp(3724549076.000003 s since 1904-01-01), "数值 2"=-40.9000015258789}, {"数值"=timestamp(3724549176.000003 s since 1904-01-01), "数值 2"=-40.7999992370605}, {"数值"=timestamp(3724549276.000003 s since 1904-01-01), "数值 2"=-39.5}, {"数值"=timestamp(3724549376.000003 s since 1904-01-01), "数值 2"=-38.5999984741211}, {"数值"=timestamp(3724549476.000003 s since 1904-01-01), "数值 2"=-39.9000015258789}, {"数值"=timestamp(3724549576.000003 s since 1904-01-01), "数值 2"=-41.0}, {"数值"=timestamp(3724549676.000003 s since 1904-01-01), "数值 2"=-41.0}, {"数值"=timestamp(3724549776.000003 s since 1904-01-01), "数值 2"=-39.7000007629395}, {"数值"=timestamp(3724549876.000003 s since 1904-01-01), "数值 2"=-38.5999984741211}, {"数值"=timestamp(3724549976.000003 s since 1904-01-01), "数值 2"=67.5}, {"数值"=timestamp(3724550076.000003 s since 1904-01-01), "数值 2"=85.3000030517578}, {"数值"=timestamp(3724550176.000003 s since 1904-01-01), "数值 2"=85.0999984741211}, {"数值"=timestamp(3724550276.000003 s since 1904-01-01), "数值 2"=85.0}, {"数值"=timestamp(3724550376.000003 s since 1904-01-01), "数值 2"=84.9000015258789}, {"数值"=timestamp(3724550476.000003 s since 1904-01-01), "数值 2"=84.9000015258789}, {"数值"=timestamp(3724550576.000003 s since 1904-01-01), "数值 2"=85.0}, {"数值"=timestamp(3724550676.000003 s since 1904-01-01), "数值 2"=85.0}, {"数值"=timestamp(3724550776.000003 s since 1904-01-01), "数值 2"=85.0}, {"数值"=timestamp(3724550876.000003 s since 1904-01-01), "数值 2"=85.0}, {"数值"=timestamp(3724550976.000003 s since 1904-01-01), "数值 2"=85.0}, {"数值"=timestamp(3724551076.000003 s since 1904-01-01), "数值 2"=85.0}, {"数值"=timestamp(3724551176.000003 s since 1904-01-01), "数值 2"=84.9000015258789}, {"数值"=timestamp(3724551276.000003 s since 1904-01-01), "数值 2"=85.0}, {"数值"=timestamp(3724551376.000003 s since 1904-01-01), "数值 2"=85.0}, {"数值"=timestamp(3724551476.000003 s since 1904-01-01), "数值 2"=84.9000015258789}, {"数值"=timestamp(3724551576.000003 s since 1904-01-01), "数值 2"=85.0}, {"数值"=timestamp(3724551676.000003 s since 1904-01-01), "数值 2"=85.0}, {"数值"=timestamp(3724551776.000003 s since 1904-01-01), "数值 2"=-11.1000003814697}, {"数值"=timestamp(3724551876.000003 s since 1904-01-01), "数值 2"=-41.7999992370605}, {"数值"=timestamp(3724551976.000003 s since 1904-01-01), "数值 2"=-40.5999984741211}, {"数值"=timestamp(3724552076.000003 s since 1904-01-01), "数值 2"=-40.2000007629395}, {"数值"=timestamp(3724552176.000003 s since 1904-01-01), "数值 2"=-38.0}, {"数值"=timestamp(3724552276.000003 s since 1904-01-01), "数值 2"=-38.5}, {"数值"=timestamp(3724552376.000003 s since 1904-01-01), "数值 2"=-39.4000015258789}, {"数值"=timestamp(3724552476.000003 s since 1904-01-01), "数值 2"=-40.5999984741211}, {"数值"=timestamp(3724552576.000003 s since 1904-01-01), "数值 2"=-41.2000007629395}, {"数值"=timestamp(3724552676.000003 s since 1904-01-01), "数值 2"=-40.7999992370605}, {"数值"=timestamp(3724552776.000003 s since 1904-01-01), "数值 2"=-39.4000015258789}, {"数值"=timestamp(3724552876.000003 s since 1904-01-01), "数值 2"=-38.7000007629395}, {"数值"=timestamp(3724552976.000003 s since 1904-01-01), "数值 2"=-40.0}, {"数值"=timestamp(3724553076.000003 s since 1904-01-01), "数值 2"=-41.0}, {"数值"=timestamp(3724553176.000003 s since 1904-01-01), "数值 2"=-41.0}, {"数值"=timestamp(3724553276.000003 s since 1904-01-01), "数值 2"=-40.0}, {"数值"=timestamp(3724553376.000003 s since 1904-01-01), "数值 2"=-38.5999984741211}, {"数值"=timestamp(3724553476.000003 s since 1904-01-01), "数值 2"=-39.2000007629395}, {"数值"=timestamp(3724553576.000003 s since 1904-01-01), "数值 2"=-40.7000007629395}, {"数值"=timestamp(3724553676.000003 s since 1904-01-01), "数值 2"=-41.2000007629395}, {"数值"=timestamp(3724553776.000003 s since 1904-01-01), "数值 2"=-40.7000007629395}, {"数值"=timestamp(3724553876.000003 s since 1904-01-01), "数值 2"=-39.0999984741211}, {"数值"=timestamp(3724553976.000003 s since 1904-01-01), "数值 2"=-38.7000007629395}, {"数值"=timestamp(3724554076.000003 s since 1904-01-01), "数值 2"=-39.9000015258789}, {"数值"=timestamp(3724554176.000003 s since 1904-01-01), "数值 2"=-41.0}, {"数值"=timestamp(3724554276.000003 s since 1904-01-01), "数值 2"=-41.2000007629395}, {"数值"=timestamp(3724554376.000003 s since 1904-01-01), "数值 2"=-40.0999984741211}, {"数值"=timestamp(3724554476.000003 s since 1904-01-01), "数值 2"=79.3000030517578}, {"数值"=timestamp(3724554576.000003 s since 1904-01-01), "数值 2"=86.0999984741211}, {"数值"=timestamp(3724554676.000003 s since 1904-01-01), "数值 2"=85.0999984741211}, {"数值"=timestamp(3724554776.000003 s since 1904-01-01), "数值 2"=85.0}, {"数值"=timestamp(3724554876.000003 s since 1904-01-01), "数值 2"=85.0999984741211}, {"数值"=timestamp(3724554976.000003 s since 1904-01-01), "数值 2"=84.9000015258789}, {"数值"=timestamp(3724555076.000003 s since 1904-01-01), "数值 2"=85.0999984741211}, {"数值"=timestamp(3724555176.000003 s since 1904-01-01), "数值 2"=85.0}, {"数值"=timestamp(3724555276.000003 s since 1904-01-01), "数值 2"=85.0}, {"数值"=timestamp(3724555376.000003 s since 1904-01-01), "数值 2"=85.0999984741211}, {"数值"=timestamp(3724555476.000003 s since 1904-01-01), "数值 2"=85.0}, {"数值"=timestamp(3724555576.000003 s since 1904-01-01), "数值 2"=85.0}, {"数值"=timestamp(3724555676.000003 s since 1904-01-01), "数值 2"=85.0}, {"数值"=timestamp(3724555776.000003 s since 1904-01-01), "数值 2"=85.0}, {"数值"=timestamp(3724555876.000003 s since 1904-01-01), "数值 2"=85.0}, {"数值"=timestamp(3724555976.000003 s since 1904-01-01), "数值 2"=85.0999984741211}, {"数值"=timestamp(3724556076.000003 s since 1904-01-01), "数值 2"=85.0}, {"数值"=timestamp(3724556176.000003 s since 1904-01-01), "数值 2"=84.9000015258789}, {"数值"=timestamp(3724556276.000003 s since 1904-01-01), "数值 2"=-21.5}, {"数值"=timestamp(3724556376.000003 s since 1904-01-01), "数值 2"=-42.4000015258789}, {"数值"=timestamp(3724556476.000003 s since 1904-01-01), "数值 2"=-40.5999984741211}, {"数值"=timestamp(3724556576.000003 s since 1904-01-01), "数值 2"=-40.0999984741211}, {"数值"=timestamp(3724556676.000003 s since 1904-01-01), "数值 2"=-38.0}, {"数值"=timestamp(3724556776.000003 s since 1904-01-01), "数值 2"=-38.5}, {"数值"=timestamp(3724556876.000003 s since 1904-01-01), "数值 2"=-39.5999984741211}, {"数值"=timestamp(3724556976.000003 s since 1904-01-01), "数值 2"=-40.2000007629395}, {"数值"=timestamp(3724557076.000003 s since 1904-01-01), "数值 2"=-40.4000015258789}, {"数值"=timestamp(3724557176.000003 s since 1904-01-01), "数值 2"=-40.4000015258789}, {"数值"=timestamp(3724557276.000003 s since 1904-01-01), "数值 2"=-40.5}, {"数值"=timestamp(3724557376.000003 s since 1904-01-01), "数值 2"=-40.2000007629395}, {"数值"=timestamp(3724557476.000003 s since 1904-01-01), "数值 2"=-39.0}, {"数值"=timestamp(3724557576.000003 s since 1904-01-01), "数值 2"=-39.0999984741211}, {"数值"=timestamp(3724557676.000003 s since 1904-01-01), "数值 2"=-40.7999992370605}, {"数值"=timestamp(3724557776.000003 s since 1904-01-01), "数值 2"=-41.0999984741211}, {"数值"=timestamp(3724557876.000003 s since 1904-01-01), "数值 2"=-40.7000007629395}, {"数值"=timestamp(3724557976.000003 s since 1904-01-01), "数值 2"=-38.9000015258789}, {"数值"=timestamp(3724558076.000003 s since 1904-01-01), "数值 2"=-38.7000007629395}, {"数值"=timestamp(3724558176.000003 s since 1904-01-01), "数值 2"=-40.2999992370605}, {"数值"=timestamp(3724558276.000003 s since 1904-01-01), "数值 2"=-41.2000007629395}, {"数值"=timestamp(3724558376.000003 s since 1904-01-01), "数值 2"=-40.7999992370605}, {"数值"=timestamp(3724558476.000003 s since 1904-01-01), "数值 2"=-39.5999984741211}, {"数值"=timestamp(3724558576.000003 s since 1904-01-01), "数值 2"=-38.5}, {"数值"=timestamp(3724558676.000003 s since 1904-01-01), "数值 2"=-39.7999992370605}, {"数值"=timestamp(3724558776.000003 s since 1904-01-01), "数值 2"=-40.9000015258789}, {"数值"=timestamp(3724558876.000003 s since 1904-01-01), "数值 2"=-41.0999984741211}, {"数值"=timestamp(3724558976.000003 s since 1904-01-01), "数值 2"=86.6999969482422}, {"数值"=timestamp(3724559076.000003 s since 1904-01-01), "数值 2"=85.9000015258789}, {"数值"=timestamp(3724559176.000003 s since 1904-01-01), "数值 2"=85.1999969482422}, {"数值"=timestamp(3724559276.000003 s since 1904-01-01), "数值 2"=85.0}, {"数值"=timestamp(3724559376.000003 s since 1904-01-01), "数值 2"=85.0999984741211}, {"数值"=timestamp(3724559476.000003 s since 1904-01-01), "数值 2"=85.0}, {"数值"=timestamp(3724559576.000003 s since 1904-01-01), "数值 2"=85.0999984741211}, {"数值"=timestamp(3724559676.000003 s since 1904-01-01), "数值 2"=85.0999984741211}, {"数值"=timestamp(3724559776.000003 s since 1904-01-01), "数值 2"=84.9000015258789}, {"数值"=timestamp(3724559876.000003 s since 1904-01-01), "数值 2"=85.0}, {"数值"=timestamp(3724559976.000003 s since 1904-01-01), "数值 2"=85.0}, {"数值"=timestamp(3724560076.000003 s since 1904-01-01), "数值 2"=85.0999984741211}, {"数值"=timestamp(3724560176.000003 s since 1904-01-01), "数值 2"=85.0}, {"数值"=timestamp(3724560276.000003 s since 1904-01-01), "数值 2"=84.9000015258789}, {"数值"=timestamp(3724560376.000003 s since 1904-01-01), "数值 2"=85.0}, {"数值"=timestamp(3724560476.000003 s since 1904-01-01), "数值 2"=85.0}, {"数值"=timestamp(3724560576.000003 s since 1904-01-01), "数值 2"=85.0}, {"数值"=timestamp(3724560676.000003 s since 1904-01-01), "数值 2"=85.0}, {"数值"=timestamp(3724560776.000003 s since 1904-01-01), "数值 2"=-28.1000003814697}, {"数值"=timestamp(3724560876.000003 s since 1904-01-01), "数值 2"=-42.0999984741211}, {"数值"=timestamp(3724560976.000003 s since 1904-01-01), "数值 2"=-40.7999992370605}, {"数值"=timestamp(3724561076.000003 s since 1904-01-01), "数值 2"=-40.0999984741211}, {"数值"=timestamp(3724561176.000003 s since 1904-01-01), "数值 2"=-38.0}, {"数值"=timestamp(3724561276.000003 s since 1904-01-01), "数值 2"=-38.4000015258789}, {"数值"=timestamp(3724561376.000003 s since 1904-01-01), "数值 2"=-39.4000015258789}, {"数值"=timestamp(3724561476.000003 s since 1904-01-01), "数值 2"=-40.7999992370605}, {"数值"=timestamp(3724561576.000003 s since 1904-01-01), "数值 2"=-41.2000007629395}, {"数值"=timestamp(3724561676.000003 s since 1904-01-01), "数值 2"=-40.5}, {"数值"=timestamp(3724561776.000003 s since 1904-01-01), "数值 2"=-39.0}, {"数值"=timestamp(3724561876.000003 s since 1904-01-01), "数值 2"=-38.7000007629395}, {"数值"=timestamp(3724561976.000003 s since 1904-01-01), "数值 2"=-40.2000007629395}, {"数值"=timestamp(3724562076.000003 s since 1904-01-01), "数值 2"=-41.0999984741211}, {"数值"=timestamp(3724562176.000003 s since 1904-01-01), "数值 2"=-41.0999984741211}, {"数值"=timestamp(3724562276.000003 s since 1904-01-01), "数值 2"=-39.7000007629395}, {"数值"=timestamp(3724562376.000003 s since 1904-01-01), "数值 2"=-38.5999984741211}, {"数值"=timestamp(3724562476.000003 s since 1904-01-01), "数值 2"=-39.0999984741211}, {"数值"=timestamp(3724562576.000003 s since 1904-01-01), "数值 2"=-40.7999992370605}, {"数值"=timestamp(3724562676.000003 s since 1904-01-01), "数值 2"=-41.2000007629395}, {"数值"=timestamp(3724562776.000003 s since 1904-01-01), "数值 2"=-40.7000007629395}, {"数值"=timestamp(3724562876.000003 s since 1904-01-01), "数值 2"=-38.7999992370605}, {"数值"=timestamp(3724562976.000003 s since 1904-01-01), "数值 2"=-38.7000007629395}, {"数值"=timestamp(3724563076.000003 s since 1904-01-01), "数值 2"=-39.5999984741211}, {"数值"=timestamp(3724563176.000003 s since 1904-01-01), "数值 2"=-41.0}, {"数值"=timestamp(3724563276.000003 s since 1904-01-01), "数值 2"=-41.2000007629395}, {"数值"=timestamp(3724563376.000003 s since 1904-01-01), "数值 2"=-40.2000007629395}, {"数值"=timestamp(3724563476.000003 s since 1904-01-01), "数值 2"=89.8000030517578}, {"数值"=timestamp(3724563576.000003 s since 1904-01-01), "数值 2"=85.6999969482422}, {"数值"=timestamp(3724563676.000003 s since 1904-01-01), "数值 2"=85.1999969482422}, {"数值"=timestamp(3724563776.000003 s since 1904-01-01), "数值 2"=85.0}, {"数值"=timestamp(3724563876.000003 s since 1904-01-01), "数值 2"=85.0}, {"数值"=timestamp(3724563976.000003 s since 1904-01-01), "数值 2"=85.0}, {"数值"=timestamp(3724564076.000003 s since 1904-01-01), "数值 2"=85.0}, {"数值"=timestamp(3724564176.000003 s since 1904-01-01), "数值 2"=85.0}, {"数值"=timestamp(3724564276.000003 s since 1904-01-01), "数值 2"=85.0}, {"数值"=timestamp(3724564376.000003 s since 1904-01-01), "数值 2"=85.0999984741211}, {"数值"=timestamp(3724564476.000003 s since 1904-01-01), "数值 2"=85.0999984741211}, {"数值"=timestamp(3724564576.000003 s since 1904-01-01), "数值 2"=84.9000015258789}, {"数值"=timestamp(3724564676.000003 s since 1904-01-01), "数值 2"=85.0}, {"数值"=timestamp(3724564776.000003 s since 1904-01-01), "数值 2"=85.0}, {"数值"=timestamp(3724564876.000003 s since 1904-01-01), "数值 2"=85.0999984741211}, {"数值"=timestamp(3724564976.000003 s since 1904-01-01), "数值 2"=84.9000015258789}, {"数值"=timestamp(3724565076.000003 s since 1904-01-01), "数值 2"=85.0}, {"数值"=timestamp(3724565176.000003 s since 1904-01-01), "数值 2"=85.0}, {"数值"=timestamp(3724565276.000003 s since 1904-01-01), "数值 2"=-33.7999992370605}, {"数值"=timestamp(3724565376.000003 s since 1904-01-01), "数值 2"=-41.9000015258789}, {"数值"=timestamp(3724565476.000003 s since 1904-01-01), "数值 2"=-40.7000007629395}, {"数值"=timestamp(3724565576.000003 s since 1904-01-01), "数值 2"=-39.7999992370605}, {"数值"=timestamp(3724565676.000003 s since 1904-01-01), "数值 2"=-37.9000015258789}, {"数值"=timestamp(3724565776.000003 s since 1904-01-01), "数值 2"=-38.2999992370605}, {"数值"=timestamp(3724565876.000003 s since 1904-01-01), "数值 2"=-39.4000015258789}, {"数值"=timestamp(3724565976.000003 s since 1904-01-01), "数值 2"=-40.7999992370605}, {"数值"=timestamp(3724566076.000003 s since 1904-01-01), "数值 2"=-41.4000015258789}, {"数值"=timestamp(3724566176.000003 s since 1904-01-01), "数值 2"=-40.7000007629395}, {"数值"=timestamp(3724566276.000003 s since 1904-01-01), "数值 2"=-39.4000015258789}, {"数值"=timestamp(3724566376.000003 s since 1904-01-01), "数值 2"=-38.4000015258789}, {"数值"=timestamp(3724566476.000003 s since 1904-01-01), "数值 2"=-39.7999992370605}, {"数值"=timestamp(3724566576.000003 s since 1904-01-01), "数值 2"=-40.9000015258789}, {"数值"=timestamp(3724566676.000003 s since 1904-01-01), "数值 2"=-41.2000007629395}, {"数值"=timestamp(3724566776.000003 s since 1904-01-01), "数值 2"=-40.4000015258789}, {"数值"=timestamp(3724566876.000003 s since 1904-01-01), "数值 2"=-38.7000007629395}, {"数值"=timestamp(3724566976.000003 s since 1904-01-01), "数值 2"=-38.9000015258789}, {"数值"=timestamp(3724567076.000003 s since 1904-01-01), "数值 2"=-40.4000015258789}, {"数值"=timestamp(3724567176.000003 s since 1904-01-01), "数值 2"=-41.2000007629395}, {"数值"=timestamp(3724567276.000003 s since 1904-01-01), "数值 2"=-40.7999992370605}, {"数值"=timestamp(3724567376.000003 s since 1904-01-01), "数值 2"=-39.4000015258789}, {"数值"=timestamp(3724567476.000003 s since 1904-01-01), "数值 2"=-38.5999984741211}, {"数值"=timestamp(3724567576.000003 s since 1904-01-01), "数值 2"=-40.0}, {"数值"=timestamp(3724567676.000003 s since 1904-01-01), "数值 2"=-41.0}, {"数值"=timestamp(3724567776.000003 s since 1904-01-01), "数值 2"=-41.0}, {"数值"=timestamp(3724567876.000003 s since 1904-01-01), "数值 2"=-40.0}, {"数值"=timestamp(3724567976.000003 s since 1904-01-01), "数值 2"=64.1999969482422}, {"数值"=timestamp(3724568076.000003 s since 1904-01-01), "数值 2"=85.5}, {"数值"=timestamp(3724568176.000003 s since 1904-01-01), "数值 2"=85.0999984741211}, {"数值"=timestamp(3724568276.000003 s since 1904-01-01), "数值 2"=85.0999984741211}, {"数值"=timestamp(3724568376.000003 s since 1904-01-01), "数值 2"=85.0999984741211}, {"数值"=timestamp(3724568476.000003 s since 1904-01-01), "数值 2"=84.9000015258789}, {"数值"=timestamp(3724568576.000003 s since 1904-01-01), "数值 2"=85.0}, {"数值"=timestamp(3724568676.000003 s since 1904-01-01), "数值 2"=85.0}, {"数值"=timestamp(3724568776.000003 s since 1904-01-01), "数值 2"=85.0}, {"数值"=timestamp(3724568876.000003 s since 1904-01-01), "数值 2"=85.0}, {"数值"=timestamp(3724568976.000003 s since 1904-01-01), "数值 2"=85.0}, {"数值"=timestamp(3724569076.000003 s since 1904-01-01), "数值 2"=85.0}, {"数值"=timestamp(3724569176.000003 s since 1904-01-01), "数值 2"=85.0}, {"数值"=timestamp(3724569276.000003 s since 1904-01-01), "数值 2"=85.0}, {"数值"=timestamp(3724569376.000003 s since 1904-01-01), "数值 2"=85.0}, {"数值"=timestamp(3724569476.000003 s since 1904-01-01), "数值 2"=85.0999984741211}, {"数值"=timestamp(3724569576.000003 s since 1904-01-01), "数值 2"=85.0}, {"数值"=timestamp(3724569676.000003 s since 1904-01-01), "数值 2"=85.0}, {"数值"=timestamp(3724569776.000003 s since 1904-01-01), "数值 2"=-7.19999980926514}, {"数值"=timestamp(3724569876.000003 s since 1904-01-01), "数值 2"=-41.7999992370605}, {"数值"=timestamp(3724569976.000003 s since 1904-01-01), "数值 2"=-40.7000007629395}, {"数值"=timestamp(3724570076.000003 s since 1904-01-01), "数值 2"=-40.4000015258789}, {"数值"=timestamp(3724570176.000003 s since 1904-01-01), "数值 2"=-38.0}, {"数值"=timestamp(3724570276.000003 s since 1904-01-01), "数值 2"=-38.5}, {"数值"=timestamp(3724570376.000003 s since 1904-01-01), "数值 2"=-39.2999992370605}, {"数值"=timestamp(3724570476.000003 s since 1904-01-01), "数值 2"=-40.9000015258789}, {"数值"=timestamp(3724570576.000003 s since 1904-01-01), "数值 2"=-41.2000007629395}, {"数值"=timestamp(3724570676.000003 s since 1904-01-01), "数值 2"=-40.5999984741211}, {"数值"=timestamp(3724570776.000003 s since 1904-01-01), "数值 2"=-38.7000007629395}, {"数值"=timestamp(3724570876.000003 s since 1904-01-01), "数值 2"=-38.7999992370605}, {"数值"=timestamp(3724570976.000003 s since 1904-01-01), "数值 2"=-40.2999992370605}, {"数值"=timestamp(3724571076.000003 s since 1904-01-01), "数值 2"=-41.2000007629395}, {"数值"=timestamp(3724571176.000003 s since 1904-01-01), "数值 2"=-40.9000015258789}, {"数值"=timestamp(3724571276.000003 s since 1904-01-01), "数值 2"=-39.7999992370605}, {"数值"=timestamp(3724571376.000003 s since 1904-01-01), "数值 2"=-38.5999984741211}, {"数值"=timestamp(3724571476.000003 s since 1904-01-01), "数值 2"=-39.5999984741211}, {"数值"=timestamp(3724571576.000003 s since 1904-01-01), "数值 2"=-40.7000007629395}, {"数值"=timestamp(3724571676.000003 s since 1904-01-01), "数值 2"=-41.0999984741211}, {"数值"=timestamp(3724571776.000003 s since 1904-01-01), "数值 2"=-40.2999992370605}, {"数值"=timestamp(3724571876.000003 s since 1904-01-01), "数值 2"=-38.9000015258789}, {"数值"=timestamp(3724571976.000003 s since 1904-01-01), "数值 2"=-39.0}, {"数值"=timestamp(3724572076.000003 s since 1904-01-01), "数值 2"=-40.5}, {"数值"=timestamp(3724572176.000003 s since 1904-01-01), "数值 2"=-41.0999984741211}, {"数值"=timestamp(3724572276.000003 s since 1904-01-01), "数值 2"=-40.5999984741211}, {"数值"=timestamp(3724572376.000003 s since 1904-01-01), "数值 2"=-39.0999984741211}, {"数值"=timestamp(3724572476.000003 s since 1904-01-01), "数值 2"=78.3000030517578}, {"数值"=timestamp(3724572576.000003 s since 1904-01-01), "数值 2"=85.1999969482422}, {"数值"=timestamp(3724572676.000003 s since 1904-01-01), "数值 2"=85.0999984741211}, {"数值"=timestamp(3724572776.000003 s since 1904-01-01), "数值 2"=85.0}, {"数值"=timestamp(3724572876.000003 s since 1904-01-01), "数值 2"=84.9000015258789}, {"数值"=timestamp(3724572976.000003 s since 1904-01-01), "数值 2"=85.0}, {"数值"=timestamp(3724573076.000003 s since 1904-01-01), "数值 2"=85.0}, {"数值"=timestamp(3724573176.000003 s since 1904-01-01), "数值 2"=85.0}, {"数值"=timestamp(3724573276.000003 s since 1904-01-01), "数值 2"=85.0}, {"数值"=timestamp(3724573376.000003 s since 1904-01-01), "数值 2"=85.0}, {"数值"=timestamp(3724573476.000003 s since 1904-01-01), "数值 2"=85.0}, {"数值"=timestamp(3724573576.000003 s since 1904-01-01), "数值 2"=85.0999984741211}, {"数值"=timestamp(3724573676.000003 s since 1904-01-01), "数值 2"=85.0}, {"数值"=timestamp(3724573776.000003 s since 1904-01-01), "数值 2"=85.0}, {"数值"=timestamp(3724573876.000003 s since 1904-01-01), "数值 2"=85.0999984741211}, {"数值"=timestamp(3724573976.000003 s since 1904-01-01), "数值 2"=85.0999984741211}, {"数值"=timestamp(3724574076.000003 s since 1904-01-01), "数值 2"=85.0999984741211}, {"数值"=timestamp(3724574176.000003 s since 1904-01-01), "数值 2"=85.0}, {"数值"=timestamp(3724574276.000003 s since 1904-01-01), "数值 2"=-18.7000007629395}, {"数值"=timestamp(3724574376.000003 s since 1904-01-01), "数值 2"=-42.7000007629395}, {"数值"=timestamp(3724574476.000003 s since 1904-01-01), "数值 2"=-41.0}, {"数值"=timestamp(3724574576.000003 s since 1904-01-01), "数值 2"=-40.2000007629395}, {"数值"=timestamp(3724574676.000003 s since 1904-01-01), "数值 2"=-38.0}, {"数值"=timestamp(3724574776.000003 s since 1904-01-01), "数值 2"=-38.5999984741211}, {"数值"=timestamp(3724574876.000003 s since 1904-01-01), "数值 2"=-39.5999984741211}, {"数值"=timestamp(3724574976.000003 s since 1904-01-01), "数值 2"=-40.7999992370605}, {"数值"=timestamp(3724575076.000003 s since 1904-01-01), "数值 2"=-41.2000007629395}, {"数值"=timestamp(3724575176.000003 s since 1904-01-01), "数值 2"=-40.2999992370605}, {"数值"=timestamp(3724575276.000003 s since 1904-01-01), "数值 2"=-38.9000015258789}, {"数值"=timestamp(3724575376.000003 s since 1904-01-01), "数值 2"=-39.0}, {"数值"=timestamp(3724575476.000003 s since 1904-01-01), "数值 2"=-40.5999984741211}, {"数值"=timestamp(3724575576.000003 s since 1904-01-01), "数值 2"=-41.0999984741211}, {"数值"=timestamp(3724575676.000003 s since 1904-01-01), "数值 2"=-40.5999984741211}, {"数值"=timestamp(3724575776.000003 s since 1904-01-01), "数值 2"=-39.2999992370605}, {"数值"=timestamp(3724575876.000003 s since 1904-01-01), "数值 2"=-38.7000007629395}, {"数值"=timestamp(3724575976.000003 s since 1904-01-01), "数值 2"=-40.0}, {"数值"=timestamp(3724576076.000003 s since 1904-01-01), "数值 2"=-41.0}, {"数值"=timestamp(3724576176.000003 s since 1904-01-01), "数值 2"=-41.0999984741211}, {"数值"=timestamp(3724576276.000003 s since 1904-01-01), "数值 2"=-39.7999992370605}, {"数值"=timestamp(3724576376.000003 s since 1904-01-01), "数值 2"=-38.5}, {"数值"=timestamp(3724576476.000003 s since 1904-01-01), "数值 2"=-39.0999984741211}, {"数值"=timestamp(3724576576.000003 s since 1904-01-01), "数值 2"=-40.7999992370605}, {"数值"=timestamp(3724576676.000003 s since 1904-01-01), "数值 2"=-41.2000007629395}, {"数值"=timestamp(3724576776.000003 s since 1904-01-01), "数值 2"=-40.5999984741211}, {"数值"=timestamp(3724576876.000003 s since 1904-01-01), "数值 2"=-38.7000007629395}, {"数值"=timestamp(3724576976.000003 s since 1904-01-01), "数值 2"=86.1999969482422}, {"数值"=timestamp(3724577076.000003 s since 1904-01-01), "数值 2"=85.8000030517578}, {"数值"=timestamp(3724577176.000003 s since 1904-01-01), "数值 2"=85.0999984741211}, {"数值"=timestamp(3724577276.000003 s since 1904-01-01), "数值 2"=85.0}, {"数值"=timestamp(3724577376.000003 s since 1904-01-01), "数值 2"=85.0999984741211}, {"数值"=timestamp(3724577476.000003 s since 1904-01-01), "数值 2"=85.0}, {"数值"=timestamp(3724577576.000003 s since 1904-01-01), "数值 2"=85.0}, {"数值"=timestamp(3724577676.000003 s since 1904-01-01), "数值 2"=85.0}, {"数值"=timestamp(3724577776.000003 s since 1904-01-01), "数值 2"=85.0}, {"数值"=timestamp(3724577876.000003 s since 1904-01-01), "数值 2"=85.0}, {"数值"=timestamp(3724577976.000003 s since 1904-01-01), "数值 2"=85.0}, {"数值"=timestamp(3724578076.000003 s since 1904-01-01), "数值 2"=85.0}, {"数值"=timestamp(3724578176.000003 s since 1904-01-01), "数值 2"=85.0}, {"数值"=timestamp(3724578276.000003 s since 1904-01-01), "数值 2"=85.0}, {"数值"=timestamp(3724578376.000003 s since 1904-01-01), "数值 2"=85.0}, {"数值"=timestamp(3724578476.000003 s since 1904-01-01), "数值 2"=85.0}, {"数值"=timestamp(3724578576.000003 s since 1904-01-01), "数值 2"=85.0999984741211}, {"数值"=timestamp(3724578676.000003 s since 1904-01-01), "数值 2"=85.0999984741211}, {"数值"=timestamp(3724578776.000003 s since 1904-01-01), "数值 2"=-27.6000003814697}, {"数值"=timestamp(3724578876.000003 s since 1904-01-01), "数值 2"=-42.2000007629395}, {"数值"=timestamp(3724578976.000003 s since 1904-01-01), "数值 2"=-40.5}, {"数值"=timestamp(3724579076.000003 s since 1904-01-01), "数值 2"=-40.0999984741211}, {"数值"=timestamp(3724579176.000003 s since 1904-01-01), "数值 2"=-38.0}, {"数值"=timestamp(3724579276.000003 s since 1904-01-01), "数值 2"=-38.5999984741211}, {"数值"=timestamp(3724579376.000003 s since 1904-01-01), "数值 2"=-39.5}, {"数值"=timestamp(3724579476.000003 s since 1904-01-01), "数值 2"=-40.7000007629395}, {"数值"=timestamp(3724579576.000003 s since 1904-01-01), "数值 2"=-41.2000007629395}, {"数值"=timestamp(3724579676.000003 s since 1904-01-01), "数值 2"=-40.5999984741211}, {"数值"=timestamp(3724579776.000003 s since 1904-01-01), "数值 2"=-39.2000007629395}, {"数值"=timestamp(3724579876.000003 s since 1904-01-01), "数值 2"=-38.7999992370605}, {"数值"=timestamp(3724579976.000003 s since 1904-01-01), "数值 2"=-40.4000015258789}, {"数值"=timestamp(3724580076.000003 s since 1904-01-01), "数值 2"=-41.0}, {"数值"=timestamp(3724580176.000003 s since 1904-01-01), "数值 2"=-40.7000007629395}, {"数值"=timestamp(3724580276.000003 s since 1904-01-01), "数值 2"=-39.5}, {"数值"=timestamp(3724580376.000003 s since 1904-01-01), "数值 2"=-38.5999984741211}, {"数值"=timestamp(3724580476.000003 s since 1904-01-01), "数值 2"=-40.0999984741211}, {"数值"=timestamp(3724580576.000003 s since 1904-01-01), "数值 2"=-40.9000015258789}, {"数值"=timestamp(3724580676.000003 s since 1904-01-01), "数值 2"=-41.0999984741211}, {"数值"=timestamp(3724580776.000003 s since 1904-01-01), "数值 2"=-40.0}, {"数值"=timestamp(3724580876.000003 s since 1904-01-01), "数值 2"=-38.5999984741211}, {"数值"=timestamp(3724580976.000003 s since 1904-01-01), "数值 2"=-38.9000015258789}, {"数值"=timestamp(3724581076.000003 s since 1904-01-01), "数值 2"=-40.5}, {"数值"=timestamp(3724581176.000003 s since 1904-01-01), "数值 2"=-41.0999984741211}, {"数值"=timestamp(3724581276.000003 s since 1904-01-01), "数值 2"=-40.5999984741211}, {"数值"=timestamp(3724581376.000003 s since 1904-01-01), "数值 2"=-39.2000007629395}, {"数值"=timestamp(3724581476.000003 s since 1904-01-01), "数值 2"=89.9000015258789}, {"数值"=timestamp(3724581576.000003 s since 1904-01-01), "数值 2"=85.5}, {"数值"=timestamp(3724581676.000003 s since 1904-01-01), "数值 2"=85.0999984741211}, {"数值"=timestamp(3724581776.000003 s since 1904-01-01), "数值 2"=85.0}, {"数值"=timestamp(3724581876.000003 s since 1904-01-01), "数值 2"=85.0}, {"数值"=timestamp(3724581976.000003 s since 1904-01-01), "数值 2"=85.0}, {"数值"=timestamp(3724582076.000003 s since 1904-01-01), "数值 2"=85.0}, {"数值"=timestamp(3724582176.000003 s since 1904-01-01), "数值 2"=85.0}, {"数值"=timestamp(3724582276.000003 s since 1904-01-01), "数值 2"=85.0999984741211}, {"数值"=timestamp(3724582376.000003 s since 1904-01-01), "数值 2"=85.0}, {"数值"=timestamp(3724582476.000003 s since 1904-01-01), "数值 2"=84.9000015258789}, {"数值"=timestamp(3724582576.000003 s since 1904-01-01), "数值 2"=85.0}, {"数值"=timestamp(3724582676.000003 s since 1904-01-01), "数值 2"=85.0}, {"数值"=timestamp(3724582776.000003 s since 1904-01-01), "数值 2"=85.0}, {"数值"=timestamp(3724582876.000003 s since 1904-01-01), "数值 2"=85.0}, {"数值"=timestamp(3724582976.000003 s since 1904-01-01), "数值 2"=85.0}, {"数值"=timestamp(3724583076.000003 s since 1904-01-01), "数值 2"=85.0}, {"数值"=timestamp(3724583176.000003 s since 1904-01-01), "数值 2"=85.0}, {"数值"=timestamp(3724583276.000003 s since 1904-01-01), "数值 2"=-33.7000007629395}, {"数值"=timestamp(3724583376.000003 s since 1904-01-01), "数值 2"=-41.5}, {"数值"=timestamp(3724583476.000003 s since 1904-01-01), "数值 2"=-40.5}, {"数值"=timestamp(3724583576.000003 s since 1904-01-01), "数值 2"=-40.0}, {"数值"=timestamp(3724583676.000003 s since 1904-01-01), "数值 2"=-38.0}, {"数值"=timestamp(3724583776.000003 s since 1904-01-01), "数值 2"=-38.5}, {"数值"=timestamp(3724583876.000003 s since 1904-01-01), "数值 2"=-39.7999992370605}, {"数值"=timestamp(3724583976.000003 s since 1904-01-01), "数值 2"=-40.9000015258789}, {"数值"=timestamp(3724584076.000003 s since 1904-01-01), "数值 2"=-41.0999984741211}, {"数值"=timestamp(3724584176.000003 s since 1904-01-01), "数值 2"=-40.2999992370605}, {"数值"=timestamp(3724584276.000003 s since 1904-01-01), "数值 2"=-38.9000015258789}, {"数值"=timestamp(3724584376.000003 s since 1904-01-01), "数值 2"=-38.7999992370605}, {"数值"=timestamp(3724584476.000003 s since 1904-01-01), "数值 2"=-40.7000007629395}, {"数值"=timestamp(3724584576.000003 s since 1904-01-01), "数值 2"=-41.2000007629395}, {"数值"=timestamp(3724584676.000003 s since 1904-01-01), "数值 2"=-40.7999992370605}, {"数值"=timestamp(3724584776.000003 s since 1904-01-01), "数值 2"=-39.2999992370605}, {"数值"=timestamp(3724584876.000003 s since 1904-01-01), "数值 2"=-38.7000007629395}, {"数值"=timestamp(3724584976.000003 s since 1904-01-01), "数值 2"=-39.5999984741211}, {"数值"=timestamp(3724585076.000003 s since 1904-01-01), "数值 2"=-40.7999992370605}, {"数值"=timestamp(3724585176.000003 s since 1904-01-01), "数值 2"=-41.0999984741211}, {"数值"=timestamp(3724585276.000003 s since 1904-01-01), "数值 2"=-40.4000015258789}, {"数值"=timestamp(3724585376.000003 s since 1904-01-01), "数值 2"=-38.7000007629395}, {"数值"=timestamp(3724585476.000003 s since 1904-01-01), "数值 2"=-39.0999984741211}, {"数值"=timestamp(3724585576.000003 s since 1904-01-01), "数值 2"=-40.2999992370605}, {"数值"=timestamp(3724585676.000003 s since 1904-01-01), "数值 2"=-40.9000015258789}, {"数值"=timestamp(3724585776.000003 s since 1904-01-01), "数值 2"=-40.7999992370605}, {"数值"=timestamp(3724585876.000003 s since 1904-01-01), "数值 2"=-39.5}, {"数值"=timestamp(3724585976.000003 s since 1904-01-01), "数值 2"=90.8000030517578}, {"数值"=timestamp(3724586076.000003 s since 1904-01-01), "数值 2"=85.1999969482422}, {"数值"=timestamp(3724586176.000003 s since 1904-01-01), "数值 2"=85.0}, {"数值"=timestamp(3724586276.000003 s since 1904-01-01), "数值 2"=85.0}, {"数值"=timestamp(3724586376.000003 s since 1904-01-01), "数值 2"=85.0}, {"数值"=timestamp(3724586476.000003 s since 1904-01-01), "数值 2"=85.0}, {"数值"=timestamp(3724586576.000003 s since 1904-01-01), "数值 2"=85.0}, {"数值"=timestamp(3724586676.000003 s since 1904-01-01), "数值 2"=85.0999984741211}, {"数值"=timestamp(3724586776.000003 s since 1904-01-01), "数值 2"=85.0}, {"数值"=timestamp(3724586876.000003 s since 1904-01-01), "数值 2"=85.0}, {"数值"=timestamp(3724586976.000003 s since 1904-01-01), "数值 2"=85.0999984741211}, {"数值"=timestamp(3724587076.000003 s since 1904-01-01), "数值 2"=85.0999984741211}, {"数值"=timestamp(3724587176.000003 s since 1904-01-01), "数值 2"=85.0}, {"数值"=timestamp(3724587276.000003 s since 1904-01-01), "数值 2"=85.0}, {"数值"=timestamp(3724587376.000003 s since 1904-01-01), "数值 2"=85.0999984741211}, {"数值"=timestamp(3724587476.000003 s since 1904-01-01), "数值 2"=84.9000015258789}, {"数值"=timestamp(3724587576.000003 s since 1904-01-01), "数值 2"=85.0}, {"数值"=timestamp(3724587676.000003 s since 1904-01-01), "数值 2"=85.0}, {"数值"=timestamp(3724587776.000003 s since 1904-01-01), "数值 2"=-37.7999992370605}, {"数值"=timestamp(3724587876.000003 s since 1904-01-01), "数值 2"=-42.0999984741211}, {"数值"=timestamp(3724587976.000003 s since 1904-01-01), "数值 2"=-40.9000015258789}, {"数值"=timestamp(3724588076.000003 s since 1904-01-01), "数值 2"=-40.2999992370605}, {"数值"=timestamp(3724588176.000003 s since 1904-01-01), "数值 2"=-38.2000007629395}, {"数值"=timestamp(3724588276.000003 s since 1904-01-01), "数值 2"=-38.7000007629395}, {"数值"=timestamp(3724588376.000003 s since 1904-01-01), "数值 2"=-39.7000007629395}, {"数值"=timestamp(3724588476.000003 s since 1904-01-01), "数值 2"=-41.0}, {"数值"=timestamp(3724588576.000003 s since 1904-01-01), "数值 2"=-41.2000007629395}, {"数值"=timestamp(3724588676.000003 s since 1904-01-01), "数值 2"=-40.5}, {"数值"=timestamp(3724588776.000003 s since 1904-01-01), "数值 2"=-38.7000007629395}, {"数值"=timestamp(3724588876.000003 s since 1904-01-01), "数值 2"=-38.9000015258789}, {"数值"=timestamp(3724588976.000003 s since 1904-01-01), "数值 2"=-40.4000015258789}, {"数值"=timestamp(3724589076.000003 s since 1904-01-01), "数值 2"=-41.0999984741211}, {"数值"=timestamp(3724589176.000003 s since 1904-01-01), "数值 2"=-40.5999984741211}, {"数值"=timestamp(3724589276.000003 s since 1904-01-01), "数值 2"=-39.4000015258789}, {"数值"=timestamp(3724589376.000003 s since 1904-01-01), "数值 2"=-38.7000007629395}, {"数值"=timestamp(3724589476.000003 s since 1904-01-01), "数值 2"=-40.2000007629395}, {"数值"=timestamp(3724589576.000003 s since 1904-01-01), "数值 2"=-41.0}, {"数值"=timestamp(3724589676.000003 s since 1904-01-01), "数值 2"=-40.9000015258789}, {"数值"=timestamp(3724589776.000003 s since 1904-01-01), "数值 2"=-39.9000015258789}, {"数值"=timestamp(3724589876.000003 s since 1904-01-01), "数值 2"=-38.5999984741211}, {"数值"=timestamp(3724589976.000003 s since 1904-01-01), "数值 2"=-39.2999992370605}, {"数值"=timestamp(3724590076.000003 s since 1904-01-01), "数值 2"=-40.7999992370605}, {"数值"=timestamp(3724590176.000003 s since 1904-01-01), "数值 2"=-41.0999984741211}, {"数值"=timestamp(3724590276.000003 s since 1904-01-01), "数值 2"=-40.4000015258789}, {"数值"=timestamp(3724590376.000003 s since 1904-01-01), "数值 2"=-39.0999984741211}, {"数值"=timestamp(3724590476.000003 s since 1904-01-01), "数值 2"=78.4000015258789}, {"数值"=timestamp(3724590576.000003 s since 1904-01-01), "数值 2"=85.0999984741211}, {"数值"=timestamp(3724590676.000003 s since 1904-01-01), "数值 2"=85.0999984741211}, {"数值"=timestamp(3724590776.000003 s since 1904-01-01), "数值 2"=85.0999984741211}, {"数值"=timestamp(3724590876.000003 s since 1904-01-01), "数值 2"=85.0}, {"数值"=timestamp(3724590976.000003 s since 1904-01-01), "数值 2"=85.0}, {"数值"=timestamp(3724591076.000003 s since 1904-01-01), "数值 2"=85.0}, {"数值"=timestamp(3724591176.000003 s since 1904-01-01), "数值 2"=85.0999984741211}, {"数值"=timestamp(3724591276.000003 s since 1904-01-01), "数值 2"=84.9000015258789}, {"数值"=timestamp(3724591376.000003 s since 1904-01-01), "数值 2"=85.0}, {"数值"=timestamp(3724591476.000003 s since 1904-01-01), "数值 2"=85.0}, {"数值"=timestamp(3724591576.000003 s since 1904-01-01), "数值 2"=85.0999984741211}, {"数值"=timestamp(3724591676.000003 s since 1904-01-01), "数值 2"=85.0}, {"数值"=timestamp(3724591776.000003 s since 1904-01-01), "数值 2"=85.0}, {"数值"=timestamp(3724591876.000003 s since 1904-01-01), "数值 2"=84.9000015258789}, {"数值"=timestamp(3724591976.000003 s since 1904-01-01), "数值 2"=84.9000015258789}, {"数值"=timestamp(3724592076.000003 s since 1904-01-01), "数值 2"=85.0}, {"数值"=timestamp(3724592176.000003 s since 1904-01-01), "数值 2"=84.9000015258789}, {"数值"=timestamp(3724592276.000003 s since 1904-01-01), "数值 2"=-15.8999996185303}, {"数值"=timestamp(3724592376.000003 s since 1904-01-01), "数值 2"=-41.5999984741211}, {"数值"=timestamp(3724592476.000003 s since 1904-01-01), "数值 2"=-40.9000015258789}, {"数值"=timestamp(3724592576.000003 s since 1904-01-01), "数值 2"=-40.2999992370605}, {"数值"=timestamp(3724592676.000003 s since 1904-01-01), "数值 2"=-38.0999984741211}, {"数值"=timestamp(3724592776.000003 s since 1904-01-01), "数值 2"=-38.5999984741211}, {"数值"=timestamp(3724592876.000003 s since 1904-01-01), "数值 2"=-39.5999984741211}, {"数值"=timestamp(3724592976.000003 s since 1904-01-01), "数值 2"=-41.0}, {"数值"=timestamp(3724593076.000003 s since 1904-01-01), "数值 2"=-41.2000007629395}, {"数值"=timestamp(3724593176.000003 s since 1904-01-01), "数值 2"=-40.5}, {"数值"=timestamp(3724593276.000003 s since 1904-01-01), "数值 2"=-38.7000007629395}, {"数值"=timestamp(3724593376.000003 s since 1904-01-01), "数值 2"=-38.9000015258789}, {"数值"=timestamp(3724593476.000003 s since 1904-01-01), "数值 2"=-40.5}, {"数值"=timestamp(3724593576.000003 s since 1904-01-01), "数值 2"=-41.0999984741211}, {"数值"=timestamp(3724593676.000003 s since 1904-01-01), "数值 2"=-40.7000007629395}, {"数值"=timestamp(3724593776.000003 s since 1904-01-01), "数值 2"=-39.5}, {"数值"=timestamp(3724593876.000003 s since 1904-01-01), "数值 2"=-38.7000007629395}, {"数值"=timestamp(3724593976.000003 s since 1904-01-01), "数值 2"=-39.7999992370605}, {"数值"=timestamp(3724594076.000003 s since 1904-01-01), "数值 2"=-40.9000015258789}, {"数值"=timestamp(3724594176.000003 s since 1904-01-01), "数值 2"=-41.0}, {"数值"=timestamp(3724594276.000003 s since 1904-01-01), "数值 2"=-40.2000007629395}, {"数值"=timestamp(3724594376.000003 s since 1904-01-01), "数值 2"=-38.7999992370605}, {"数值"=timestamp(3724594476.000003 s since 1904-01-01), "数值 2"=-39.0}, {"数值"=timestamp(3724594576.000003 s since 1904-01-01), "数值 2"=-40.5999984741211}, {"数值"=timestamp(3724594676.000003 s since 1904-01-01), "数值 2"=-41.0}, {"数值"=timestamp(3724594776.000003 s since 1904-01-01), "数值 2"=-40.7000007629395}, {"数值"=timestamp(3724594876.000003 s since 1904-01-01), "数值 2"=-39.5999984741211}, {"数值"=timestamp(3724594976.000003 s since 1904-01-01), "数值 2"=86.0999984741211}, {"数值"=timestamp(3724595076.000003 s since 1904-01-01), "数值 2"=85.9000015258789}, {"数值"=timestamp(3724595176.000003 s since 1904-01-01), "数值 2"=85.0999984741211}, {"数值"=timestamp(3724595276.000003 s since 1904-01-01), "数值 2"=85.0}, {"数值"=timestamp(3724595376.000003 s since 1904-01-01), "数值 2"=85.0999984741211}, {"数值"=timestamp(3724595476.000003 s since 1904-01-01), "数值 2"=85.0}, {"数值"=timestamp(3724595576.000003 s since 1904-01-01), "数值 2"=85.0}, {"数值"=timestamp(3724595676.000003 s since 1904-01-01), "数值 2"=85.0}, {"数值"=timestamp(3724595776.000003 s since 1904-01-01), "数值 2"=84.9000015258789}, {"数值"=timestamp(3724595876.000003 s since 1904-01-01), "数值 2"=84.9000015258789}, {"数值"=timestamp(3724595976.000003 s since 1904-01-01), "数值 2"=85.0}, {"数值"=timestamp(3724596076.000003 s since 1904-01-01), "数值 2"=84.9000015258789}, {"数值"=timestamp(3724596176.000003 s since 1904-01-01), "数值 2"=85.0}, {"数值"=timestamp(3724596276.000003 s since 1904-01-01), "数值 2"=85.0999984741211}, {"数值"=timestamp(3724596376.000003 s since 1904-01-01), "数值 2"=84.9000015258789}, {"数值"=timestamp(3724596476.000003 s since 1904-01-01), "数值 2"=85.0}, {"数值"=timestamp(3724596576.000003 s since 1904-01-01), "数值 2"=84.9000015258789}, {"数值"=timestamp(3724596676.000003 s since 1904-01-01), "数值 2"=85.0999984741211}, {"数值"=timestamp(3724596776.000003 s since 1904-01-01), "数值 2"=-26.7000007629395}, {"数值"=timestamp(3724596876.000003 s since 1904-01-01), "数值 2"=-42.7000007629395}, {"数值"=timestamp(3724596976.000003 s since 1904-01-01), "数值 2"=-40.9000015258789}, {"数值"=timestamp(3724597076.000003 s since 1904-01-01), "数值 2"=-39.9000015258789}, {"数值"=timestamp(3724597176.000003 s since 1904-01-01), "数值 2"=-38.0999984741211}, {"数值"=timestamp(3724597276.000003 s since 1904-01-01), "数值 2"=-38.7999992370605}, {"数值"=timestamp(3724597376.000003 s since 1904-01-01), "数值 2"=-39.7000007629395}, {"数值"=timestamp(3724597476.000003 s since 1904-01-01), "数值 2"=-40.9000015258789}, {"数值"=timestamp(3724597576.000003 s since 1904-01-01), "数值 2"=-41.0999984741211}, {"数值"=timestamp(3724597676.000003 s since 1904-01-01), "数值 2"=-40.2999992370605}, {"数值"=timestamp(3724597776.000003 s since 1904-01-01), "数值 2"=-38.9000015258789}, {"数值"=timestamp(3724597876.000003 s since 1904-01-01), "数值 2"=-38.9000015258789}, {"数值"=timestamp(3724597976.000003 s since 1904-01-01), "数值 2"=-40.4000015258789}, {"数值"=timestamp(3724598076.000003 s since 1904-01-01), "数值 2"=-41.0999984741211}, {"数值"=timestamp(3724598176.000003 s since 1904-01-01), "数值 2"=-40.7000007629395}, {"数值"=timestamp(3724598276.000003 s since 1904-01-01), "数值 2"=-39.5}, {"数值"=timestamp(3724598376.000003 s since 1904-01-01), "数值 2"=-38.5999984741211}, {"数值"=timestamp(3724598476.000003 s since 1904-01-01), "数值 2"=-39.7000007629395}, {"数值"=timestamp(3724598576.000003 s since 1904-01-01), "数值 2"=-40.9000015258789}, {"数值"=timestamp(3724598676.000003 s since 1904-01-01), "数值 2"=-41.2000007629395}, {"数值"=timestamp(3724598776.000003 s since 1904-01-01), "数值 2"=-40.2000007629395}, {"数值"=timestamp(3724598876.000003 s since 1904-01-01), "数值 2"=-38.9000015258789}, {"数值"=timestamp(3724598976.000003 s since 1904-01-01), "数值 2"=-38.5999984741211}, {"数值"=timestamp(3724599076.000003 s since 1904-01-01), "数值 2"=-40.5999984741211}, {"数值"=timestamp(3724599176.000003 s since 1904-01-01), "数值 2"=-41.0}, {"数值"=timestamp(3724599276.000003 s since 1904-01-01), "数值 2"=-40.9000015258789}, {"数值"=timestamp(3724599376.000003 s since 1904-01-01), "数值 2"=-39.4000015258789}, {"数值"=timestamp(3724599476.000003 s since 1904-01-01), "数值 2"=90.4000015258789}, {"数值"=timestamp(3724599576.000003 s since 1904-01-01), "数值 2"=85.5}, {"数值"=timestamp(3724599676.000003 s since 1904-01-01), "数值 2"=85.0999984741211}, {"数值"=timestamp(3724599776.000003 s since 1904-01-01), "数值 2"=85.0999984741211}, {"数值"=timestamp(3724599876.000003 s since 1904-01-01), "数值 2"=85.0999984741211}, {"数值"=timestamp(3724599976.000003 s since 1904-01-01), "数值 2"=85.0999984741211}, {"数值"=timestamp(3724600076.000003 s since 1904-01-01), "数值 2"=84.9000015258789}, {"数值"=timestamp(3724600176.000003 s since 1904-01-01), "数值 2"=85.0}, {"数值"=timestamp(3724600276.000003 s since 1904-01-01), "数值 2"=85.0}, {"数值"=timestamp(3724600376.000003 s since 1904-01-01), "数值 2"=85.0}, {"数值"=timestamp(3724600476.000003 s since 1904-01-01), "数值 2"=85.0999984741211}, {"数值"=timestamp(3724600576.000003 s since 1904-01-01), "数值 2"=85.0}, {"数值"=timestamp(3724600676.000003 s since 1904-01-01), "数值 2"=85.0}, {"数值"=timestamp(3724600776.000003 s since 1904-01-01), "数值 2"=85.0999984741211}, {"数值"=timestamp(3724600876.000003 s since 1904-01-01), "数值 2"=84.9000015258789}, {"数值"=timestamp(3724600976.000003 s since 1904-01-01), "数值 2"=85.0}, {"数值"=timestamp(3724601076.000003 s since 1904-01-01), "数值 2"=85.0999984741211}, {"数值"=timestamp(3724601176.000003 s since 1904-01-01), "数值 2"=84.9000015258789}, {"数值"=timestamp(3724601276.000003 s since 1904-01-01), "数值 2"=-32.0999984741211}, {"数值"=timestamp(3724601376.000003 s since 1904-01-01), "数值 2"=-41.7000007629395}, {"数值"=timestamp(3724601476.000003 s since 1904-01-01), "数值 2"=-40.5}, {"数值"=timestamp(3724601576.000003 s since 1904-01-01), "数值 2"=-40.0999984741211}, {"数值"=timestamp(3724601676.000003 s since 1904-01-01), "数值 2"=-38.0}, {"数值"=timestamp(3724601776.000003 s since 1904-01-01), "数值 2"=-38.5999984741211}, {"数值"=timestamp(3724601876.000003 s since 1904-01-01), "数值 2"=-39.5999984741211}, {"数值"=timestamp(3724601976.000003 s since 1904-01-01), "数值 2"=-40.7999992370605}, {"数值"=timestamp(3724602076.000003 s since 1904-01-01), "数值 2"=-41.0999984741211}, {"数值"=timestamp(3724602176.000003 s since 1904-01-01), "数值 2"=-40.5}, {"数值"=timestamp(3724602276.000003 s since 1904-01-01), "数值 2"=-38.9000015258789}, {"数值"=timestamp(3724602376.000003 s since 1904-01-01), "数值 2"=-38.7000007629395}, {"数值"=timestamp(3724602476.000003 s since 1904-01-01), "数值 2"=-40.5999984741211}, {"数值"=timestamp(3724602576.000003 s since 1904-01-01), "数值 2"=-41.0}, {"数值"=timestamp(3724602676.000003 s since 1904-01-01), "数值 2"=-40.9000015258789}, {"数值"=timestamp(3724602776.000003 s since 1904-01-01), "数值 2"=-39.5}, {"数值"=timestamp(3724602876.000003 s since 1904-01-01), "数值 2"=-38.5}, {"数值"=timestamp(3724602976.000003 s since 1904-01-01), "数值 2"=-39.0999984741211}, {"数值"=timestamp(3724603076.000003 s since 1904-01-01), "数值 2"=-40.9000015258789}, {"数值"=timestamp(3724603176.000003 s since 1904-01-01), "数值 2"=-41.0999984741211}, {"数值"=timestamp(3724603276.000003 s since 1904-01-01), "数值 2"=-40.5}, {"数值"=timestamp(3724603376.000003 s since 1904-01-01), "数值 2"=-38.7000007629395}, {"数值"=timestamp(3724603476.000003 s since 1904-01-01), "数值 2"=-38.9000015258789}, {"数值"=timestamp(3724603576.000003 s since 1904-01-01), "数值 2"=-40.5}, {"数值"=timestamp(3724603676.000003 s since 1904-01-01), "数值 2"=-41.2000007629395}, {"数值"=timestamp(3724603776.000003 s since 1904-01-01), "数值 2"=-40.7999992370605}, {"数值"=timestamp(3724603876.000003 s since 1904-01-01), "数值 2"=-39.5}, {"数值"=timestamp(3724603976.000003 s since 1904-01-01), "数值 2"=90.5999984741211}, {"数值"=timestamp(3724604076.000003 s since 1904-01-01), "数值 2"=85.1999969482422}, {"数值"=timestamp(3724604176.000003 s since 1904-01-01), "数值 2"=85.0}, {"数值"=timestamp(3724604276.000003 s since 1904-01-01), "数值 2"=85.0}, {"数值"=timestamp(3724604376.000003 s since 1904-01-01), "数值 2"=85.0}, {"数值"=timestamp(3724604476.000003 s since 1904-01-01), "数值 2"=85.0}, {"数值"=timestamp(3724604576.000003 s since 1904-01-01), "数值 2"=85.0}, {"数值"=timestamp(3724604676.000003 s since 1904-01-01), "数值 2"=85.0}, {"数值"=timestamp(3724604776.000003 s since 1904-01-01), "数值 2"=85.0}, {"数值"=timestamp(3724604876.000003 s since 1904-01-01), "数值 2"=85.0999984741211}, {"数值"=timestamp(3724604976.000003 s since 1904-01-01), "数值 2"=84.9000015258789}, {"数值"=timestamp(3724605076.000003 s since 1904-01-01), "数值 2"=85.0999984741211}, {"数值"=timestamp(3724605176.000003 s since 1904-01-01), "数值 2"=84.9000015258789}, {"数值"=timestamp(3724605276.000003 s since 1904-01-01), "数值 2"=85.0}, {"数值"=timestamp(3724605376.000003 s since 1904-01-01), "数值 2"=85.0}, {"数值"=timestamp(3724605476.000003 s since 1904-01-01), "数值 2"=85.0}, {"数值"=timestamp(3724605576.000003 s since 1904-01-01), "数值 2"=85.0}, {"数值"=timestamp(3724605676.000003 s since 1904-01-01), "数值 2"=85.0999984741211}, {"数值"=timestamp(3724605776.000003 s since 1904-01-01), "数值 2"=-36.7999992370605}, {"数值"=timestamp(3724605876.000003 s since 1904-01-01), "数值 2"=-41.5999984741211}, {"数值"=timestamp(3724605976.000003 s since 1904-01-01), "数值 2"=-40.7000007629395}, {"数值"=timestamp(3724606076.000003 s since 1904-01-01), "数值 2"=-40.0}, {"数值"=timestamp(3724606176.000003 s since 1904-01-01), "数值 2"=-38.0}, {"数值"=timestamp(3724606276.000003 s since 1904-01-01), "数值 2"=-38.5}, {"数值"=timestamp(3724606376.000003 s since 1904-01-01), "数值 2"=-39.5999984741211}, {"数值"=timestamp(3724606476.000003 s since 1904-01-01), "数值 2"=-41.0}, {"数值"=timestamp(3724606576.000003 s since 1904-01-01), "数值 2"=-41.2000007629395}, {"数值"=timestamp(3724606676.000003 s since 1904-01-01), "数值 2"=-40.2999992370605}, {"数值"=timestamp(3724606776.000003 s since 1904-01-01), "数值 2"=-38.9000015258789}, {"数值"=timestamp(3724606876.000003 s since 1904-01-01), "数值 2"=-38.7999992370605}, {"数值"=timestamp(3724606976.000003 s since 1904-01-01), "数值 2"=-40.5999984741211}, {"数值"=timestamp(3724607076.000003 s since 1904-01-01), "数值 2"=-41.0}, {"数值"=timestamp(3724607176.000003 s since 1904-01-01), "数值 2"=-40.9000015258789}, {"数值"=timestamp(3724607276.000003 s since 1904-01-01), "数值 2"=-39.2999992370605}, {"数值"=timestamp(3724607376.000003 s since 1904-01-01), "数值 2"=-38.5999984741211}, {"数值"=timestamp(3724607476.000003 s since 1904-01-01), "数值 2"=-39.7999992370605}, {"数值"=timestamp(3724607576.000003 s since 1904-01-01), "数值 2"=-41.0}, {"数值"=timestamp(3724607676.000003 s since 1904-01-01), "数值 2"=-41.0999984741211}, {"数值"=timestamp(3724607776.000003 s since 1904-01-01), "数值 2"=-40.2000007629395}, {"数值"=timestamp(3724607876.000003 s since 1904-01-01), "数值 2"=-38.5}, {"数值"=timestamp(3724607976.000003 s since 1904-01-01), "数值 2"=-39.0}, {"数值"=timestamp(3724608076.000003 s since 1904-01-01), "数值 2"=-40.5999984741211}, {"数值"=timestamp(3724608176.000003 s since 1904-01-01), "数值 2"=-41.2000007629395}, {"数值"=timestamp(3724608276.000003 s since 1904-01-01), "数值 2"=-40.5999984741211}, {"数值"=timestamp(3724608376.000003 s since 1904-01-01), "数值 2"=-39.2999992370605}, {"数值"=timestamp(3724608476.000003 s since 1904-01-01), "数值 2"=89.0}, {"数值"=timestamp(3724608576.000003 s since 1904-01-01), "数值 2"=85.0999984741211}, {"数值"=timestamp(3724608676.000003 s since 1904-01-01), "数值 2"=85.0999984741211}, {"数值"=timestamp(3724608776.000003 s since 1904-01-01), "数值 2"=85.0}, {"数值"=timestamp(3724608876.000003 s since 1904-01-01), "数值 2"=85.0}, {"数值"=timestamp(3724608976.000003 s since 1904-01-01), "数值 2"=85.0}, {"数值"=timestamp(3724609076.000003 s since 1904-01-01), "数值 2"=85.0}, {"数值"=timestamp(3724609176.000003 s since 1904-01-01), "数值 2"=85.0}, {"数值"=timestamp(3724609276.000003 s since 1904-01-01), "数值 2"=85.0}, {"数值"=timestamp(3724609376.000003 s since 1904-01-01), "数值 2"=85.0}, {"数值"=timestamp(3724609476.000003 s since 1904-01-01), "数值 2"=85.0}, {"数值"=timestamp(3724609576.000003 s since 1904-01-01), "数值 2"=85.0}, {"数值"=timestamp(3724609676.000003 s since 1904-01-01), "数值 2"=85.0}, {"数值"=timestamp(3724609776.000003 s since 1904-01-01), "数值 2"=85.0}, {"数值"=timestamp(3724609876.000003 s since 1904-01-01), "数值 2"=84.9000015258789}, {"数值"=timestamp(3724609976.000003 s since 1904-01-01), "数值 2"=84.9000015258789}, {"数值"=timestamp(3724610076.000003 s since 1904-01-01), "数值 2"=84.9000015258789}, {"数值"=timestamp(3724610176.000003 s since 1904-01-01), "数值 2"=84.9000015258789}, {"数值"=timestamp(3724610276.000003 s since 1904-01-01), "数值 2"=-15.1000003814697}, {"数值"=timestamp(3724610376.000003 s since 1904-01-01), "数值 2"=-42.4000015258789}, {"数值"=timestamp(3724610476.000003 s since 1904-01-01), "数值 2"=-40.9000015258789}, {"数值"=timestamp(3724610576.000003 s since 1904-01-01), "数值 2"=-39.5}, {"数值"=timestamp(3724610676.000003 s since 1904-01-01), "数值 2"=-38.2000007629395}, {"数值"=timestamp(3724610776.000003 s since 1904-01-01), "数值 2"=-38.7999992370605}, {"数值"=timestamp(3724610876.000003 s since 1904-01-01), "数值 2"=-39.7000007629395}, {"数值"=timestamp(3724610976.000003 s since 1904-01-01), "数值 2"=-40.9000015258789}, {"数值"=timestamp(3724611076.000003 s since 1904-01-01), "数值 2"=-41.0999984741211}, {"数值"=timestamp(3724611176.000003 s since 1904-01-01), "数值 2"=-40.4000015258789}, {"数值"=timestamp(3724611276.000003 s since 1904-01-01), "数值 2"=-38.5999984741211}, {"数值"=timestamp(3724611376.000003 s since 1904-01-01), "数值 2"=-39.2000007629395}, {"数值"=timestamp(3724611476.000003 s since 1904-01-01), "数值 2"=-40.7000007629395}, {"数值"=timestamp(3724611576.000003 s since 1904-01-01), "数值 2"=-41.0999984741211}, {"数值"=timestamp(3724611676.000003 s since 1904-01-01), "数值 2"=-40.5999984741211}, {"数值"=timestamp(3724611776.000003 s since 1904-01-01), "数值 2"=-39.0999984741211}, {"数值"=timestamp(3724611876.000003 s since 1904-01-01), "数值 2"=-38.7999992370605}, {"数值"=timestamp(3724611976.000003 s since 1904-01-01), "数值 2"=-40.2999992370605}, {"数值"=timestamp(3724612076.000003 s since 1904-01-01), "数值 2"=-41.0}, {"数值"=timestamp(3724612176.000003 s since 1904-01-01), "数值 2"=-40.9000015258789}, {"数值"=timestamp(3724612276.000003 s since 1904-01-01), "数值 2"=-39.5999984741211}, {"数值"=timestamp(3724612376.000003 s since 1904-01-01), "数值 2"=-38.5999984741211}, {"数值"=timestamp(3724612476.000003 s since 1904-01-01), "数值 2"=-39.7999992370605}, {"数值"=timestamp(3724612576.000003 s since 1904-01-01), "数值 2"=-40.9000015258789}, {"数值"=timestamp(3724612676.000003 s since 1904-01-01), "数值 2"=-41.0999984741211}, {"数值"=timestamp(3724612776.000003 s since 1904-01-01), "数值 2"=-40.0}, {"数值"=timestamp(3724612876.000003 s since 1904-01-01), "数值 2"=-38.5999984741211}, {"数值"=timestamp(3724612976.000003 s since 1904-01-01), "数值 2"=83.3000030517578}, {"数值"=timestamp(3724613076.000003 s since 1904-01-01), "数值 2"=85.4000015258789}, {"数值"=timestamp(3724613176.000003 s since 1904-01-01), "数值 2"=85.1999969482422}, {"数值"=timestamp(3724613276.000003 s since 1904-01-01), "数值 2"=85.0999984741211}, {"数值"=timestamp(3724613376.000003 s since 1904-01-01), "数值 2"=85.0}, {"数值"=timestamp(3724613476.000003 s since 1904-01-01), "数值 2"=85.0}, {"数值"=timestamp(3724613576.000003 s since 1904-01-01), "数值 2"=85.0}, {"数值"=timestamp(3724613676.000003 s since 1904-01-01), "数值 2"=85.0}, {"数值"=timestamp(3724613776.000003 s since 1904-01-01), "数值 2"=85.0}, {"数值"=timestamp(3724613876.000003 s since 1904-01-01), "数值 2"=85.0}, {"数值"=timestamp(3724613976.000003 s since 1904-01-01), "数值 2"=85.0999984741211}, {"数值"=timestamp(3724614076.000003 s since 1904-01-01), "数值 2"=85.0}, {"数值"=timestamp(3724614176.000003 s since 1904-01-01), "数值 2"=85.0}, {"数值"=timestamp(3724614276.000003 s since 1904-01-01), "数值 2"=85.0}, {"数值"=timestamp(3724614376.000003 s since 1904-01-01), "数值 2"=85.0}, {"数值"=timestamp(3724614476.000003 s since 1904-01-01), "数值 2"=85.0}, {"数值"=timestamp(3724614576.000003 s since 1904-01-01), "数值 2"=85.0}, {"数值"=timestamp(3724614676.000003 s since 1904-01-01), "数值 2"=85.0999984741211}, {"数值"=timestamp(3724614776.000003 s since 1904-01-01), "数值 2"=-25.1000003814697}, {"数值"=timestamp(3724614876.000003 s since 1904-01-01), "数值 2"=-42.2999992370605}, {"数值"=timestamp(3724614976.000003 s since 1904-01-01), "数值 2"=-40.9000015258789}, {"数值"=timestamp(3724615076.000003 s since 1904-01-01), "数值 2"=-39.7999992370605}, {"数值"=timestamp(3724615176.000003 s since 1904-01-01), "数值 2"=-38.0999984741211}, {"数值"=timestamp(3724615276.000003 s since 1904-01-01), "数值 2"=-38.7000007629395}, {"数值"=timestamp(3724615376.000003 s since 1904-01-01), "数值 2"=-39.7000007629395}, {"数值"=timestamp(3724615476.000003 s since 1904-01-01), "数值 2"=-41.0}, {"数值"=timestamp(3724615576.000003 s since 1904-01-01), "数值 2"=-41.0}, {"数值"=timestamp(3724615676.000003 s since 1904-01-01), "数值 2"=-40.2999992370605}, {"数值"=timestamp(3724615776.000003 s since 1904-01-01), "数值 2"=-38.5999984741211}, {"数值"=timestamp(3724615876.000003 s since 1904-01-01), "数值 2"=-39.5}, {"数值"=timestamp(3724615976.000003 s since 1904-01-01), "数值 2"=-40.5999984741211}, {"数值"=timestamp(3724616076.000003 s since 1904-01-01), "数值 2"=-41.0999984741211}, {"数值"=timestamp(3724616176.000003 s since 1904-01-01), "数值 2"=-40.5}, {"数值"=timestamp(3724616276.000003 s since 1904-01-01), "数值 2"=-39.0}, {"数值"=timestamp(3724616376.000003 s since 1904-01-01), "数值 2"=-38.5999984741211}, {"数值"=timestamp(3724616476.000003 s since 1904-01-01), "数值 2"=-40.5}, {"数值"=timestamp(3724616576.000003 s since 1904-01-01), "数值 2"=-41.0}, {"数值"=timestamp(3724616676.000003 s since 1904-01-01), "数值 2"=-40.9000015258789}, {"数值"=timestamp(3724616776.000003 s since 1904-01-01), "数值 2"=-39.4000015258789}, {"数值"=timestamp(3724616876.000003 s since 1904-01-01), "数值 2"=-38.7000007629395}, {"数值"=timestamp(3724616976.000003 s since 1904-01-01), "数值 2"=-39.5999984741211}, {"数值"=timestamp(3724617076.000003 s since 1904-01-01), "数值 2"=-40.9000015258789}, {"数值"=timestamp(3724617176.000003 s since 1904-01-01), "数值 2"=-40.9000015258789}, {"数值"=timestamp(3724617276.000003 s since 1904-01-01), "数值 2"=-40.0999984741211}, {"数值"=timestamp(3724617376.000003 s since 1904-01-01), "数值 2"=-38.7000007629395}, {"数值"=timestamp(3724617476.000003 s since 1904-01-01), "数值 2"=89.1999969482422}, {"数值"=timestamp(3724617576.000003 s since 1904-01-01), "数值 2"=85.5999984741211}, {"数值"=timestamp(3724617676.000003 s since 1904-01-01), "数值 2"=85.0999984741211}, {"数值"=timestamp(3724617776.000003 s since 1904-01-01), "数值 2"=85.0}, {"数值"=timestamp(3724617876.000003 s since 1904-01-01), "数值 2"=85.0999984741211}, {"数值"=timestamp(3724617976.000003 s since 1904-01-01), "数值 2"=85.0999984741211}, {"数值"=timestamp(3724618076.000003 s since 1904-01-01), "数值 2"=85.0}, {"数值"=timestamp(3724618176.000003 s since 1904-01-01), "数值 2"=85.0}, {"数值"=timestamp(3724618276.000003 s since 1904-01-01), "数值 2"=85.0}, {"数值"=timestamp(3724618376.000003 s since 1904-01-01), "数值 2"=85.0}, {"数值"=timestamp(3724618476.000003 s since 1904-01-01), "数值 2"=85.0}, {"数值"=timestamp(3724618576.000003 s since 1904-01-01), "数值 2"=85.0}, {"数值"=timestamp(3724618676.000003 s since 1904-01-01), "数值 2"=85.0999984741211}, {"数值"=timestamp(3724618776.000003 s since 1904-01-01), "数值 2"=85.0999984741211}, {"数值"=timestamp(3724618876.000003 s since 1904-01-01), "数值 2"=84.9000015258789}, {"数值"=timestamp(3724618976.000003 s since 1904-01-01), "数值 2"=85.0}, {"数值"=timestamp(3724619076.000003 s since 1904-01-01), "数值 2"=85.0999984741211}, {"数值"=timestamp(3724619176.000003 s since 1904-01-01), "数值 2"=84.9000015258789}, {"数值"=timestamp(3724619276.000003 s since 1904-01-01), "数值 2"=-31.5}, {"数值"=timestamp(3724619376.000003 s since 1904-01-01), "数值 2"=-41.5999984741211}, {"数值"=timestamp(3724619476.000003 s since 1904-01-01), "数值 2"=-40.5999984741211}, {"数值"=timestamp(3724619576.000003 s since 1904-01-01), "数值 2"=-40.2999992370605}, {"数值"=timestamp(3724619676.000003 s since 1904-01-01), "数值 2"=-38.0}, {"数值"=timestamp(3724619776.000003 s since 1904-01-01), "数值 2"=-38.5}, {"数值"=timestamp(3724619876.000003 s since 1904-01-01), "数值 2"=-39.4000015258789}, {"数值"=timestamp(3724619976.000003 s since 1904-01-01), "数值 2"=-40.7000007629395}, {"数值"=timestamp(3724620076.000003 s since 1904-01-01), "数值 2"=-41.2999992370605}, {"数值"=timestamp(3724620176.000003 s since 1904-01-01), "数值 2"=-40.5999984741211}, {"数值"=timestamp(3724620276.000003 s since 1904-01-01), "数值 2"=-39.2000007629395}, {"数值"=timestamp(3724620376.000003 s since 1904-01-01), "数值 2"=-38.7999992370605}, {"数值"=timestamp(3724620476.000003 s since 1904-01-01), "数值 2"=-40.0999984741211}, {"数值"=timestamp(3724620576.000003 s since 1904-01-01), "数值 2"=-41.0}, {"数值"=timestamp(3724620676.000003 s since 1904-01-01), "数值 2"=-41.0}, {"数值"=timestamp(3724620776.000003 s since 1904-01-01), "数值 2"=-40.0}, {"数值"=timestamp(3724620876.000003 s since 1904-01-01), "数值 2"=-38.5999984741211}, {"数值"=timestamp(3724620976.000003 s since 1904-01-01), "数值 2"=-39.2000007629395}, {"数值"=timestamp(3724621076.000003 s since 1904-01-01), "数值 2"=-40.7000007629395}, {"数值"=timestamp(3724621176.000003 s since 1904-01-01), "数值 2"=-41.2000007629395}, {"数值"=timestamp(3724621276.000003 s since 1904-01-01), "数值 2"=-40.5}, {"数值"=timestamp(3724621376.000003 s since 1904-01-01), "数值 2"=-39.0999984741211}, {"数值"=timestamp(3724621476.000003 s since 1904-01-01), "数值 2"=-38.5999984741211}, {"数值"=timestamp(3724621576.000003 s since 1904-01-01), "数值 2"=-40.4000015258789}, {"数值"=timestamp(3724621676.000003 s since 1904-01-01), "数值 2"=-41.2000007629395}, {"数值"=timestamp(3724621776.000003 s since 1904-01-01), "数值 2"=-41.0}, {"数值"=timestamp(3724621876.000003 s since 1904-01-01), "数值 2"=-39.4000015258789}, {"数值"=timestamp(3724621976.000003 s since 1904-01-01), "数值 2"=90.5}, {"数值"=timestamp(3724622076.000003 s since 1904-01-01), "数值 2"=85.4000015258789}, {"数值"=timestamp(3724622176.000003 s since 1904-01-01), "数值 2"=85.0}, {"数值"=timestamp(3724622276.000003 s since 1904-01-01), "数值 2"=85.0999984741211}, {"数值"=timestamp(3724622376.000003 s since 1904-01-01), "数值 2"=84.9000015258789}, {"数值"=timestamp(3724622476.000003 s since 1904-01-01), "数值 2"=85.0}, {"数值"=timestamp(3724622576.000003 s since 1904-01-01), "数值 2"=85.0}, {"数值"=timestamp(3724622676.000003 s since 1904-01-01), "数值 2"=85.0}, {"数值"=timestamp(3724622776.000003 s since 1904-01-01), "数值 2"=85.0}, {"数值"=timestamp(3724622876.000003 s since 1904-01-01), "数值 2"=85.0}, {"数值"=timestamp(3724622976.000003 s since 1904-01-01), "数值 2"=85.0999984741211}, {"数值"=timestamp(3724623076.000003 s since 1904-01-01), "数值 2"=85.0}, {"数值"=timestamp(3724623176.000003 s since 1904-01-01), "数值 2"=85.0}, {"数值"=timestamp(3724623276.000003 s since 1904-01-01), "数值 2"=85.0}, {"数值"=timestamp(3724623376.000003 s since 1904-01-01), "数值 2"=85.0999984741211}, {"数值"=timestamp(3724623476.000003 s since 1904-01-01), "数值 2"=84.9000015258789}, {"数值"=timestamp(3724623576.000003 s since 1904-01-01), "数值 2"=85.0}, {"数值"=timestamp(3724623676.000003 s since 1904-01-01), "数值 2"=85.0}, {"数值"=timestamp(3724623776.000003 s since 1904-01-01), "数值 2"=-35.7999992370605}, {"数值"=timestamp(3724623876.000003 s since 1904-01-01), "数值 2"=-42.0}, {"数值"=timestamp(3724623976.000003 s since 1904-01-01), "数值 2"=-40.9000015258789}, {"数值"=timestamp(3724624076.000003 s since 1904-01-01), "数值 2"=-39.7000007629395}, {"数值"=timestamp(3724624176.000003 s since 1904-01-01), "数值 2"=-37.9000015258789}, {"数值"=timestamp(3724624276.000003 s since 1904-01-01), "数值 2"=-38.4000015258789}, {"数值"=timestamp(3724624376.000003 s since 1904-01-01), "数值 2"=-39.9000015258789}, {"数值"=timestamp(3724624476.000003 s since 1904-01-01), "数值 2"=-40.9000015258789}, {"数值"=timestamp(3724624576.000003 s since 1904-01-01), "数值 2"=-41.0999984741211}, {"数值"=timestamp(3724624676.000003 s since 1904-01-01), "数值 2"=-40.0}, {"数值"=timestamp(3724624776.000003 s since 1904-01-01), "数值 2"=-38.7000007629395}, {"数值"=timestamp(3724624876.000003 s since 1904-01-01), "数值 2"=-39.0}, {"数值"=timestamp(3724624976.000003 s since 1904-01-01), "数值 2"=-40.7000007629395}, {"数值"=timestamp(3724625076.000003 s since 1904-01-01), "数值 2"=-41.0999984741211}, {"数值"=timestamp(3724625176.000003 s since 1904-01-01), "数值 2"=-40.7000007629395}, {"数值"=timestamp(3724625276.000003 s since 1904-01-01), "数值 2"=-38.7999992370605}, {"数值"=timestamp(3724625376.000003 s since 1904-01-01), "数值 2"=-38.7999992370605}, {"数值"=timestamp(3724625476.000003 s since 1904-01-01), "数值 2"=-40.2999992370605}, {"数值"=timestamp(3724625576.000003 s since 1904-01-01), "数值 2"=-41.0}, {"数值"=timestamp(3724625676.000003 s since 1904-01-01), "数值 2"=-40.7999992370605}, {"数值"=timestamp(3724625776.000003 s since 1904-01-01), "数值 2"=-39.5999984741211}, {"数值"=timestamp(3724625876.000003 s since 1904-01-01), "数值 2"=-38.7000007629395}, {"数值"=timestamp(3724625976.000003 s since 1904-01-01), "数值 2"=-40.0999984741211}, {"数值"=timestamp(3724626076.000003 s since 1904-01-01), "数值 2"=-40.9000015258789}, {"数值"=timestamp(3724626176.000003 s since 1904-01-01), "数值 2"=-41.0}, {"数值"=timestamp(3724626276.000003 s since 1904-01-01), "数值 2"=-39.9000015258789}, {"数值"=timestamp(3724626376.000003 s since 1904-01-01), "数值 2"=-38.5999984741211}, {"数值"=timestamp(3724626476.000003 s since 1904-01-01), "数值 2"=89.3000030517578}, {"数值"=timestamp(3724626576.000003 s since 1904-01-01), "数值 2"=85.1999969482422}, {"数值"=timestamp(3724626676.000003 s since 1904-01-01), "数值 2"=85.0}, {"数值"=timestamp(3724626776.000003 s since 1904-01-01), "数值 2"=85.0}, {"数值"=timestamp(3724626876.000003 s since 1904-01-01), "数值 2"=85.0999984741211}, {"数值"=timestamp(3724626976.000003 s since 1904-01-01), "数值 2"=85.0}, {"数值"=timestamp(3724627076.000003 s since 1904-01-01), "数值 2"=85.0}, {"数值"=timestamp(3724627176.000003 s since 1904-01-01), "数值 2"=85.0}, {"数值"=timestamp(3724627276.000003 s since 1904-01-01), "数值 2"=85.0}, {"数值"=timestamp(3724627376.000003 s since 1904-01-01), "数值 2"=85.0999984741211}, {"数值"=timestamp(3724627476.000003 s since 1904-01-01), "数值 2"=84.9000015258789}, {"数值"=timestamp(3724627576.000003 s since 1904-01-01), "数值 2"=84.9000015258789}, {"数值"=timestamp(3724627676.000003 s since 1904-01-01), "数值 2"=85.0999984741211}, {"数值"=timestamp(3724627776.000003 s since 1904-01-01), "数值 2"=85.0999984741211}, {"数值"=timestamp(3724627876.000003 s since 1904-01-01), "数值 2"=85.0}, {"数值"=timestamp(3724627976.000003 s since 1904-01-01), "数值 2"=85.0999984741211}, {"数值"=timestamp(3724628076.000003 s since 1904-01-01), "数值 2"=85.0999984741211}, {"数值"=timestamp(3724628176.000003 s since 1904-01-01), "数值 2"=85.0}, {"数值"=timestamp(3724628276.000003 s since 1904-01-01), "数值 2"=-39.7999992370605}, {"数值"=timestamp(3724628376.000003 s since 1904-01-01), "数值 2"=-42.2999992370605}, {"数值"=timestamp(3724628476.000003 s since 1904-01-01), "数值 2"=-41.0}, {"数值"=timestamp(3724628576.000003 s since 1904-01-01), "数值 2"=-39.5}, {"数值"=timestamp(3724628676.000003 s since 1904-01-01), "数值 2"=-38.2000007629395}, {"数值"=timestamp(3724628776.000003 s since 1904-01-01), "数值 2"=-38.7000007629395}, {"数值"=timestamp(3724628876.000003 s since 1904-01-01), "数值 2"=-39.9000015258789}, {"数值"=timestamp(3724628976.000003 s since 1904-01-01), "数值 2"=-41.0}, {"数值"=timestamp(3724629076.000003 s since 1904-01-01), "数值 2"=-41.0999984741211}, {"数值"=timestamp(3724629176.000003 s since 1904-01-01), "数值 2"=-40.2000007629395}, {"数值"=timestamp(3724629276.000003 s since 1904-01-01), "数值 2"=-38.7000007629395}, {"数值"=timestamp(3724629376.000003 s since 1904-01-01), "数值 2"=-38.7000007629395}, {"数值"=timestamp(3724629476.000003 s since 1904-01-01), "数值 2"=-40.7000007629395}, {"数值"=timestamp(3724629576.000003 s since 1904-01-01), "数值 2"=-41.0999984741211}, {"数值"=timestamp(3724629676.000003 s since 1904-01-01), "数值 2"=-40.7999992370605}, {"数值"=timestamp(3724629776.000003 s since 1904-01-01), "数值 2"=-39.0999984741211}, {"数值"=timestamp(3724629876.000003 s since 1904-01-01), "数值 2"=-38.7000007629395}, {"数值"=timestamp(3724629976.000003 s since 1904-01-01), "数值 2"=-40.0}, {"数值"=timestamp(3724630076.000003 s since 1904-01-01), "数值 2"=-41.0}, {"数值"=timestamp(3724630176.000003 s since 1904-01-01), "数值 2"=-40.7999992370605}, {"数值"=timestamp(3724630276.000003 s since 1904-01-01), "数值 2"=-39.7999992370605}, {"数值"=timestamp(3724630376.000003 s since 1904-01-01), "数值 2"=-38.7000007629395}, {"数值"=timestamp(3724630476.000003 s since 1904-01-01), "数值 2"=-39.5999984741211}, {"数值"=timestamp(3724630576.000003 s since 1904-01-01), "数值 2"=-40.9000015258789}, {"数值"=timestamp(3724630676.000003 s since 1904-01-01), "数值 2"=-41.0999984741211}, {"数值"=timestamp(3724630776.000003 s since 1904-01-01), "数值 2"=-40.0999984741211}, {"数值"=timestamp(3724630876.000003 s since 1904-01-01), "数值 2"=-38.7000007629395}, {"数值"=timestamp(3724630976.000003 s since 1904-01-01), "数值 2"=83.0999984741211}, {"数值"=timestamp(3724631076.000003 s since 1904-01-01), "数值 2"=85.0999984741211}, {"数值"=timestamp(3724631176.000003 s since 1904-01-01), "数值 2"=85.0999984741211}, {"数值"=timestamp(3724631276.000003 s since 1904-01-01), "数值 2"=85.0}, {"数值"=timestamp(3724631376.000003 s since 1904-01-01), "数值 2"=85.0999984741211}, {"数值"=timestamp(3724631476.000003 s since 1904-01-01), "数值 2"=84.9000015258789}, {"数值"=timestamp(3724631576.000003 s since 1904-01-01), "数值 2"=85.0}, {"数值"=timestamp(3724631676.000003 s since 1904-01-01), "数值 2"=85.0}, {"数值"=timestamp(3724631776.000003 s since 1904-01-01), "数值 2"=85.0}, {"数值"=timestamp(3724631876.000003 s since 1904-01-01), "数值 2"=85.0}, {"数值"=timestamp(3724631976.000003 s since 1904-01-01), "数值 2"=85.0}, {"数值"=timestamp(3724632076.000003 s since 1904-01-01), "数值 2"=85.0}, {"数值"=timestamp(3724632176.000003 s since 1904-01-01), "数值 2"=85.0}, {"数值"=timestamp(3724632276.000003 s since 1904-01-01), "数值 2"=85.0}, {"数值"=timestamp(3724632376.000003 s since 1904-01-01), "数值 2"=85.0}, {"数值"=timestamp(3724632476.000003 s since 1904-01-01), "数值 2"=85.0}, {"数值"=timestamp(3724632576.000003 s since 1904-01-01), "数值 2"=85.0}, {"数值"=timestamp(3724632676.000003 s since 1904-01-01), "数值 2"=84.9000015258789}, {"数值"=timestamp(3724632776.000003 s since 1904-01-01), "数值 2"=-23.7000007629395}, {"数值"=timestamp(3724632876.000003 s since 1904-01-01), "数值 2"=-41.9000015258789}, {"数值"=timestamp(3724632976.000003 s since 1904-01-01), "数值 2"=-41.0}, {"数值"=timestamp(3724633076.000003 s since 1904-01-01), "数值 2"=-39.7000007629395}, {"数值"=timestamp(3724633176.000003 s since 1904-01-01), "数值 2"=-38.2000007629395}, {"数值"=timestamp(3724633276.000003 s since 1904-01-01), "数值 2"=-38.5999984741211}, {"数值"=timestamp(3724633376.000003 s since 1904-01-01), "数值 2"=-39.5}, {"数值"=timestamp(3724633476.000003 s since 1904-01-01), "数值 2"=-41.0}, {"数值"=timestamp(3724633576.000003 s since 1904-01-01), "数值 2"=-41.0999984741211}, {"数值"=timestamp(3724633676.000003 s since 1904-01-01), "数值 2"=-40.2999992370605}, {"数值"=timestamp(3724633776.000003 s since 1904-01-01), "数值 2"=-38.7000007629395}, {"数值"=timestamp(3724633876.000003 s since 1904-01-01), "数值 2"=-39.2999992370605}, {"数值"=timestamp(3724633976.000003 s since 1904-01-01), "数值 2"=-40.7000007629395}, {"数值"=timestamp(3724634076.000003 s since 1904-01-01), "数值 2"=-41.0999984741211}, {"数值"=timestamp(3724634176.000003 s since 1904-01-01), "数值 2"=-40.2999992370605}, {"数值"=timestamp(3724634276.000003 s since 1904-01-01), "数值 2"=-38.7999992370605}, {"数值"=timestamp(3724634376.000003 s since 1904-01-01), "数值 2"=-39.0}, {"数值"=timestamp(3724634476.000003 s since 1904-01-01), "数值 2"=-40.5999984741211}, {"数值"=timestamp(3724634576.000003 s since 1904-01-01), "数值 2"=-41.0999984741211}, {"数值"=timestamp(3724634676.000003 s since 1904-01-01), "数值 2"=-40.5}, {"数值"=timestamp(3724634776.000003 s since 1904-01-01), "数值 2"=-39.0}, {"数值"=timestamp(3724634876.000003 s since 1904-01-01), "数值 2"=-38.5999984741211}, {"数值"=timestamp(3724634976.000003 s since 1904-01-01), "数值 2"=-40.4000015258789}, {"数值"=timestamp(3724635076.000003 s since 1904-01-01), "数值 2"=-41.0999984741211}, {"数值"=timestamp(3724635176.000003 s since 1904-01-01), "数值 2"=-41.0}, {"数值"=timestamp(3724635276.000003 s since 1904-01-01), "数值 2"=-39.2999992370605}, {"数值"=timestamp(3724635376.000003 s since 1904-01-01), "数值 2"=-38.5999984741211}, {"数值"=timestamp(3724635476.000003 s since 1904-01-01), "数值 2"=87.9000015258789}, {"数值"=timestamp(3724635576.000003 s since 1904-01-01), "数值 2"=85.4000015258789}, {"数值"=timestamp(3724635676.000003 s since 1904-01-01), "数值 2"=85.1999969482422}, {"数值"=timestamp(3724635776.000003 s since 1904-01-01), "数值 2"=85.0}, {"数值"=timestamp(3724635876.000003 s since 1904-01-01), "数值 2"=85.0}, {"数值"=timestamp(3724635976.000003 s since 1904-01-01), "数值 2"=84.9000015258789}, {"数值"=timestamp(3724636076.000003 s since 1904-01-01), "数值 2"=85.0}, {"数值"=timestamp(3724636176.000003 s since 1904-01-01), "数值 2"=85.0999984741211}, {"数值"=timestamp(3724636276.000003 s since 1904-01-01), "数值 2"=85.0}, {"数值"=timestamp(3724636376.000003 s since 1904-01-01), "数值 2"=85.0}, {"数值"=timestamp(3724636476.000003 s since 1904-01-01), "数值 2"=85.0}, {"数值"=timestamp(3724636576.000003 s since 1904-01-01), "数值 2"=85.0}, {"数值"=timestamp(3724636676.000003 s since 1904-01-01), "数值 2"=85.0}, {"数值"=timestamp(3724636776.000003 s since 1904-01-01), "数值 2"=85.0}, {"数值"=timestamp(3724636876.000003 s since 1904-01-01), "数值 2"=85.0}, {"数值"=timestamp(3724636976.000003 s since 1904-01-01), "数值 2"=85.0}, {"数值"=timestamp(3724637076.000003 s since 1904-01-01), "数值 2"=85.0999984741211}, {"数值"=timestamp(3724637176.000003 s since 1904-01-01), "数值 2"=85.0}, {"数值"=timestamp(3724637276.000003 s since 1904-01-01), "数值 2"=-29.7999992370605}, {"数值"=timestamp(3724637376.000003 s since 1904-01-01), "数值 2"=-41.5}, {"数值"=timestamp(3724637476.000003 s since 1904-01-01), "数值 2"=-40.5}, {"数值"=timestamp(3724637576.000003 s since 1904-01-01), "数值 2"=-39.5999984741211}, {"数值"=timestamp(3724637676.000003 s since 1904-01-01), "数值 2"=-37.7000007629395}, {"数值"=timestamp(3724637776.000003 s since 1904-01-01), "数值 2"=-38.5999984741211}, {"数值"=timestamp(3724637876.000003 s since 1904-01-01), "数值 2"=-39.7000007629395}, {"数值"=timestamp(3724637976.000003 s since 1904-01-01), "数值 2"=-40.7000007629395}, {"数值"=timestamp(3724638076.000003 s since 1904-01-01), "数值 2"=-41.0}, {"数值"=timestamp(3724638176.000003 s since 1904-01-01), "数值 2"=-40.2999992370605}, {"数值"=timestamp(3724638276.000003 s since 1904-01-01), "数值 2"=-38.7999992370605}, {"数值"=timestamp(3724638376.000003 s since 1904-01-01), "数值 2"=-39.0999984741211}, {"数值"=timestamp(3724638476.000003 s since 1904-01-01), "数值 2"=-40.5999984741211}, {"数值"=timestamp(3724638576.000003 s since 1904-01-01), "数值 2"=-41.2000007629395}, {"数值"=timestamp(3724638676.000003 s since 1904-01-01), "数值 2"=-40.7000007629395}, {"数值"=timestamp(3724638776.000003 s since 1904-01-01), "数值 2"=-39.4000015258789}, {"数值"=timestamp(3724638876.000003 s since 1904-01-01), "数值 2"=-38.5999984741211}, {"数值"=timestamp(3724638976.000003 s since 1904-01-01), "数值 2"=-39.7999992370605}, {"数值"=timestamp(3724639076.000003 s since 1904-01-01), "数值 2"=-41.0}, {"数值"=timestamp(3724639176.000003 s since 1904-01-01), "数值 2"=-41.0999984741211}, {"数值"=timestamp(3724639276.000003 s since 1904-01-01), "数值 2"=-39.7999992370605}, {"数值"=timestamp(3724639376.000003 s since 1904-01-01), "数值 2"=-38.5999984741211}, {"数值"=timestamp(3724639476.000003 s since 1904-01-01), "数值 2"=-39.0999984741211}, {"数值"=timestamp(3724639576.000003 s since 1904-01-01), "数值 2"=-40.7999992370605}, {"数值"=timestamp(3724639676.000003 s since 1904-01-01), "数值 2"=-41.0999984741211}, {"数值"=timestamp(3724639776.000003 s since 1904-01-01), "数值 2"=-40.5}, {"数值"=timestamp(3724639876.000003 s since 1904-01-01), "数值 2"=-38.5999984741211}, {"数值"=timestamp(3724639976.000003 s since 1904-01-01), "数值 2"=90.0999984741211}, {"数值"=timestamp(3724640076.000003 s since 1904-01-01), "数值 2"=85.6999969482422}, {"数值"=timestamp(3724640176.000003 s since 1904-01-01), "数值 2"=85.0999984741211}, {"数值"=timestamp(3724640276.000003 s since 1904-01-01), "数值 2"=85.0999984741211}, {"数值"=timestamp(3724640376.000003 s since 1904-01-01), "数值 2"=85.0}, {"数值"=timestamp(3724640476.000003 s since 1904-01-01), "数值 2"=84.9000015258789}, {"数值"=timestamp(3724640576.000003 s since 1904-01-01), "数值 2"=85.0999984741211}, {"数值"=timestamp(3724640676.000003 s since 1904-01-01), "数值 2"=85.0}, {"数值"=timestamp(3724640776.000003 s since 1904-01-01), "数值 2"=85.0}, {"数值"=timestamp(3724640876.000003 s since 1904-01-01), "数值 2"=85.0}, {"数值"=timestamp(3724640976.000003 s since 1904-01-01), "数值 2"=85.0}, {"数值"=timestamp(3724641076.000003 s since 1904-01-01), "数值 2"=85.0}, {"数值"=timestamp(3724641176.000003 s since 1904-01-01), "数值 2"=85.0}, {"数值"=timestamp(3724641276.000003 s since 1904-01-01), "数值 2"=84.9000015258789}, {"数值"=timestamp(3724641376.000003 s since 1904-01-01), "数值 2"=85.0}, {"数值"=timestamp(3724641476.000003 s since 1904-01-01), "数值 2"=85.0}, {"数值"=timestamp(3724641576.000003 s since 1904-01-01), "数值 2"=85.0}, {"数值"=timestamp(3724641676.000003 s since 1904-01-01), "数值 2"=85.0}, {"数值"=timestamp(3724641776.000003 s since 1904-01-01), "数值 2"=-35.0}, {"数值"=timestamp(3724641876.000003 s since 1904-01-01), "数值 2"=-42.4000015258789}, {"数值"=timestamp(3724641976.000003 s since 1904-01-01), "数值 2"=-40.9000015258789}, {"数值"=timestamp(3724642076.000003 s since 1904-01-01), "数值 2"=-39.9000015258789}, {"数值"=timestamp(3724642176.000003 s since 1904-01-01), "数值 2"=-38.0}, {"数值"=timestamp(3724642276.000003 s since 1904-01-01), "数值 2"=-38.9000015258789}, {"数值"=timestamp(3724642376.000003 s since 1904-01-01), "数值 2"=-39.9000015258789}, {"数值"=timestamp(3724642476.000003 s since 1904-01-01), "数值 2"=-40.9000015258789}, {"数值"=timestamp(3724642576.000003 s since 1904-01-01), "数值 2"=-41.0}, {"数值"=timestamp(3724642676.000003 s since 1904-01-01), "数值 2"=-40.2000007629395}, {"数值"=timestamp(3724642776.000003 s since 1904-01-01), "数值 2"=-38.7000007629395}, {"数值"=timestamp(3724642876.000003 s since 1904-01-01), "数值 2"=-39.5}, {"数值"=timestamp(3724642976.000003 s since 1904-01-01), "数值 2"=-40.7999992370605}, {"数值"=timestamp(3724643076.000003 s since 1904-01-01), "数值 2"=-41.2000007629395}, {"数值"=timestamp(3724643176.000003 s since 1904-01-01), "数值 2"=-40.2999992370605}, {"数值"=timestamp(3724643276.000003 s since 1904-01-01), "数值 2"=-38.7999992370605}, {"数值"=timestamp(3724643376.000003 s since 1904-01-01), "数值 2"=-38.7999992370605}, {"数值"=timestamp(3724643476.000003 s since 1904-01-01), "数值 2"=-40.2999992370605}, {"数值"=timestamp(3724643576.000003 s since 1904-01-01), "数值 2"=-41.2000007629395}, {"数值"=timestamp(3724643676.000003 s since 1904-01-01), "数值 2"=-41.2000007629395}, {"数值"=timestamp(3724643776.000003 s since 1904-01-01), "数值 2"=-39.7999992370605}, {"数值"=timestamp(3724643876.000003 s since 1904-01-01), "数值 2"=-38.5}, {"数值"=timestamp(3724643976.000003 s since 1904-01-01), "数值 2"=-38.9000015258789}, {"数值"=timestamp(3724644076.000003 s since 1904-01-01), "数值 2"=-40.7000007629395}, {"数值"=timestamp(3724644176.000003 s since 1904-01-01), "数值 2"=-41.0999984741211}, {"数值"=timestamp(3724644276.000003 s since 1904-01-01), "数值 2"=-40.7000007629395}, {"数值"=timestamp(3724644376.000003 s since 1904-01-01), "数值 2"=-38.7999992370605}, {"数值"=timestamp(3724644476.000003 s since 1904-01-01), "数值 2"=88.9000015258789}, {"数值"=timestamp(3724644576.000003 s since 1904-01-01), "数值 2"=85.4000015258789}, {"数值"=timestamp(3724644676.000003 s since 1904-01-01), "数值 2"=85.0999984741211}, {"数值"=timestamp(3724644776.000003 s since 1904-01-01), "数值 2"=85.0999984741211}, {"数值"=timestamp(3724644876.000003 s since 1904-01-01), "数值 2"=84.9000015258789}, {"数值"=timestamp(3724644976.000003 s since 1904-01-01), "数值 2"=84.9000015258789}, {"数值"=timestamp(3724645076.000003 s since 1904-01-01), "数值 2"=85.0}, {"数值"=timestamp(3724645176.000003 s since 1904-01-01), "数值 2"=85.0}, {"数值"=timestamp(3724645276.000003 s since 1904-01-01), "数值 2"=85.0}, {"数值"=timestamp(3724645376.000003 s since 1904-01-01), "数值 2"=85.0}, {"数值"=timestamp(3724645476.000003 s since 1904-01-01), "数值 2"=85.0}, {"数值"=timestamp(3724645576.000003 s since 1904-01-01), "数值 2"=85.0}, {"数值"=timestamp(3724645676.000003 s since 1904-01-01), "数值 2"=85.0}, {"数值"=timestamp(3724645776.000003 s since 1904-01-01), "数值 2"=85.0}, {"数值"=timestamp(3724645876.000003 s since 1904-01-01), "数值 2"=85.0999984741211}, {"数值"=timestamp(3724645976.000003 s since 1904-01-01), "数值 2"=85.0}, {"数值"=timestamp(3724646076.000003 s since 1904-01-01), "数值 2"=84.9000015258789}, {"数值"=timestamp(3724646176.000003 s since 1904-01-01), "数值 2"=85.0}, {"数值"=timestamp(3724646276.000003 s since 1904-01-01), "数值 2"=-39.7000007629395}, {"数值"=timestamp(3724646376.000003 s since 1904-01-01), "数值 2"=-42.4000015258789}, {"数值"=timestamp(3724646476.000003 s since 1904-01-01), "数值 2"=-41.0}, {"数值"=timestamp(3724646576.000003 s since 1904-01-01), "数值 2"=-39.0999984741211}, {"数值"=timestamp(3724646676.000003 s since 1904-01-01), "数值 2"=-38.0}, {"数值"=timestamp(3724646776.000003 s since 1904-01-01), "数值 2"=-38.7000007629395}, {"数值"=timestamp(3724646876.000003 s since 1904-01-01), "数值 2"=-39.7999992370605}, {"数值"=timestamp(3724646976.000003 s since 1904-01-01), "数值 2"=-41.0999984741211}, {"数值"=timestamp(3724647076.000003 s since 1904-01-01), "数值 2"=-41.2000007629395}, {"数值"=timestamp(3724647176.000003 s since 1904-01-01), "数值 2"=-40.0}, {"数值"=timestamp(3724647276.000003 s since 1904-01-01), "数值 2"=-38.7000007629395}, {"数值"=timestamp(3724647376.000003 s since 1904-01-01), "数值 2"=-39.0999984741211}, {"数值"=timestamp(3724647476.000003 s since 1904-01-01), "数值 2"=-40.7999992370605}, {"数值"=timestamp(3724647576.000003 s since 1904-01-01), "数值 2"=-41.2000007629395}, {"数值"=timestamp(3724647676.000003 s since 1904-01-01), "数值 2"=-40.7000007629395}, {"数值"=timestamp(3724647776.000003 s since 1904-01-01), "数值 2"=-38.7999992370605}, {"数值"=timestamp(3724647876.000003 s since 1904-01-01), "数值 2"=-38.7000007629395}, {"数值"=timestamp(3724647976.000003 s since 1904-01-01), "数值 2"=-40.0}, {"数值"=timestamp(3724648076.000003 s since 1904-01-01), "数值 2"=-41.2000007629395}, {"数值"=timestamp(3724648176.000003 s since 1904-01-01), "数值 2"=-41.0}, {"数值"=timestamp(3724648276.000003 s since 1904-01-01), "数值 2"=-39.5999984741211}, {"数值"=timestamp(3724648376.000003 s since 1904-01-01), "数值 2"=-38.7000007629395}, {"数值"=timestamp(3724648476.000003 s since 1904-01-01), "数值 2"=-39.7999992370605}, {"数值"=timestamp(3724648576.000003 s since 1904-01-01), "数值 2"=-40.7999992370605}, {"数值"=timestamp(3724648676.000003 s since 1904-01-01), "数值 2"=-41.0999984741211}, {"数值"=timestamp(3724648776.000003 s since 1904-01-01), "数值 2"=-40.2000007629395}, {"数值"=timestamp(3724648876.000003 s since 1904-01-01), "数值 2"=-38.7999992370605}, {"数值"=timestamp(3724648976.000003 s since 1904-01-01), "数值 2"=87.0999984741211}, {"数值"=timestamp(3724649076.000003 s since 1904-01-01), "数值 2"=85.4000015258789}, {"数值"=timestamp(3724649176.000003 s since 1904-01-01), "数值 2"=85.1999969482422}, {"数值"=timestamp(3724649276.000003 s since 1904-01-01), "数值 2"=85.0}, {"数值"=timestamp(3724649376.000003 s since 1904-01-01), "数值 2"=85.0999984741211}, {"数值"=timestamp(3724649476.000003 s since 1904-01-01), "数值 2"=85.0}, {"数值"=timestamp(3724649576.000003 s since 1904-01-01), "数值 2"=85.0999984741211}, {"数值"=timestamp(3724649676.000003 s since 1904-01-01), "数值 2"=85.0999984741211}, {"数值"=timestamp(3724649776.000003 s since 1904-01-01), "数值 2"=85.0}, {"数值"=timestamp(3724649876.000003 s since 1904-01-01), "数值 2"=85.0}, {"数值"=timestamp(3724649976.000003 s since 1904-01-01), "数值 2"=85.0}, {"数值"=timestamp(3724650076.000003 s since 1904-01-01), "数值 2"=85.0}, {"数值"=timestamp(3724650176.000003 s since 1904-01-01), "数值 2"=85.0}, {"数值"=timestamp(3724650276.000003 s since 1904-01-01), "数值 2"=85.0}, {"数值"=timestamp(3724650376.000003 s since 1904-01-01), "数值 2"=85.0}, {"数值"=timestamp(3724650476.000003 s since 1904-01-01), "数值 2"=85.0}, {"数值"=timestamp(3724650576.000003 s since 1904-01-01), "数值 2"=85.0999984741211}, {"数值"=timestamp(3724650676.000003 s since 1904-01-01), "数值 2"=85.0999984741211}, {"数值"=timestamp(3724650776.000003 s since 1904-01-01), "数值 2"=-40.9000015258789}, {"数值"=timestamp(3724650876.000003 s since 1904-01-01), "数值 2"=-41.4000015258789}, {"数值"=timestamp(3724650976.000003 s since 1904-01-01), "数值 2"=-40.5999984741211}, {"数值"=timestamp(3724651076.000003 s since 1904-01-01), "数值 2"=-40.0}, {"数值"=timestamp(3724651176.000003 s since 1904-01-01), "数值 2"=-37.7999992370605}, {"数值"=timestamp(3724651276.000003 s since 1904-01-01), "数值 2"=-38.2999992370605}, {"数值"=timestamp(3724651376.000003 s since 1904-01-01), "数值 2"=-39.9000015258789}, {"数值"=timestamp(3724651476.000003 s since 1904-01-01), "数值 2"=-41.0}, {"数值"=timestamp(3724651576.000003 s since 1904-01-01), "数值 2"=-41.0}, {"数值"=timestamp(3724651676.000003 s since 1904-01-01), "数值 2"=-40.0}, {"数值"=timestamp(3724651776.000003 s since 1904-01-01), "数值 2"=-38.7000007629395}, {"数值"=timestamp(3724651876.000003 s since 1904-01-01), "数值 2"=-39.0}, {"数值"=timestamp(3724651976.000003 s since 1904-01-01), "数值 2"=-40.4000015258789}, {"数值"=timestamp(3724652076.000003 s since 1904-01-01), "数值 2"=-41.2000007629395}, {"数值"=timestamp(3724652176.000003 s since 1904-01-01), "数值 2"=-40.7999992370605}, {"数值"=timestamp(3724652276.000003 s since 1904-01-01), "数值 2"=-39.4000015258789}, {"数值"=timestamp(3724652376.000003 s since 1904-01-01), "数值 2"=-38.7000007629395}, {"数值"=timestamp(3724652476.000003 s since 1904-01-01), "数值 2"=-40.0}, {"数值"=timestamp(3724652576.000003 s since 1904-01-01), "数值 2"=-41.0}, {"数值"=timestamp(3724652676.000003 s since 1904-01-01), "数值 2"=-41.0}, {"数值"=timestamp(3724652776.000003 s since 1904-01-01), "数值 2"=-40.0}, {"数值"=timestamp(3724652876.000003 s since 1904-01-01), "数值 2"=-38.5999984741211}, {"数值"=timestamp(3724652976.000003 s since 1904-01-01), "数值 2"=-39.2000007629395}, {"数值"=timestamp(3724653076.000003 s since 1904-01-01), "数值 2"=-40.5999984741211}, {"数值"=timestamp(3724653176.000003 s since 1904-01-01), "数值 2"=-41.2000007629395}, {"数值"=timestamp(3724653276.000003 s since 1904-01-01), "数值 2"=-40.5}, {"数值"=timestamp(3724653376.000003 s since 1904-01-01), "数值 2"=-39.0}, {"数值"=timestamp(3724653476.000003 s since 1904-01-01), "数值 2"=88.4000015258789}, {"数值"=timestamp(3724653576.000003 s since 1904-01-01), "数值 2"=85.4000015258789}, {"数值"=timestamp(3724653676.000003 s since 1904-01-01), "数值 2"=85.0999984741211}, {"数值"=timestamp(3724653776.000003 s since 1904-01-01), "数值 2"=85.0}, {"数值"=timestamp(3724653876.000003 s since 1904-01-01), "数值 2"=85.0}, {"数值"=timestamp(3724653976.000003 s since 1904-01-01), "数值 2"=85.0}, {"数值"=timestamp(3724654076.000003 s since 1904-01-01), "数值 2"=85.0}, {"数值"=timestamp(3724654176.000003 s since 1904-01-01), "数值 2"=85.0}, {"数值"=timestamp(3724654276.000003 s since 1904-01-01), "数值 2"=85.0999984741211}, {"数值"=timestamp(3724654376.000003 s since 1904-01-01), "数值 2"=85.0}, {"数值"=timestamp(3724654476.000003 s since 1904-01-01), "数值 2"=85.0}, {"数值"=timestamp(3724654576.000003 s since 1904-01-01), "数值 2"=85.0}, {"数值"=timestamp(3724654676.000003 s since 1904-01-01), "数值 2"=84.9000015258789}, {"数值"=timestamp(3724654776.000003 s since 1904-01-01), "数值 2"=85.0}, {"数值"=timestamp(3724654876.000003 s since 1904-01-01), "数值 2"=84.9000015258789}, {"数值"=timestamp(3724654976.000003 s since 1904-01-01), "数值 2"=85.0}, {"数值"=timestamp(3724655076.000003 s since 1904-01-01), "数值 2"=85.0999984741211}, {"数值"=timestamp(3724655176.000003 s since 1904-01-01), "数值 2"=85.0}, {"数值"=timestamp(3724655276.000003 s since 1904-01-01), "数值 2"=-32.2000007629395}, {"数值"=timestamp(3724655376.000003 s since 1904-01-01), "数值 2"=-41.7000007629395}, {"数值"=timestamp(3724655476.000003 s since 1904-01-01), "数值 2"=-40.7999992370605}, {"数值"=timestamp(3724655576.000003 s since 1904-01-01), "数值 2"=-39.7000007629395}, {"数值"=timestamp(3724655676.000003 s since 1904-01-01), "数值 2"=-38.0}, {"数值"=timestamp(3724655776.000003 s since 1904-01-01), "数值 2"=-38.7999992370605}, {"数值"=timestamp(3724655876.000003 s since 1904-01-01), "数值 2"=-39.7999992370605}, {"数值"=timestamp(3724655976.000003 s since 1904-01-01), "数值 2"=-41.2000007629395}, {"数值"=timestamp(3724656076.000003 s since 1904-01-01), "数值 2"=-41.0}, {"数值"=timestamp(3724656176.000003 s since 1904-01-01), "数值 2"=-40.0999984741211}, {"数值"=timestamp(3724656276.000003 s since 1904-01-01), "数值 2"=-38.7000007629395}, {"数值"=timestamp(3724656376.000003 s since 1904-01-01), "数值 2"=-39.4000015258789}, {"数值"=timestamp(3724656476.000003 s since 1904-01-01), "数值 2"=-40.7999992370605}, {"数值"=timestamp(3724656576.000003 s since 1904-01-01), "数值 2"=-41.0}, {"数值"=timestamp(3724656676.000003 s since 1904-01-01), "数值 2"=-40.4000015258789}, {"数值"=timestamp(3724656776.000003 s since 1904-01-01), "数值 2"=-38.9000015258789}, {"数值"=timestamp(3724656876.000003 s since 1904-01-01), "数值 2"=-39.0999984741211}, {"数值"=timestamp(3724656976.000003 s since 1904-01-01), "数值 2"=-40.7000007629395}, {"数值"=timestamp(3724657076.000003 s since 1904-01-01), "数值 2"=-41.0}, {"数值"=timestamp(3724657176.000003 s since 1904-01-01), "数值 2"=-40.4000015258789}, {"数值"=timestamp(3724657276.000003 s since 1904-01-01), "数值 2"=-38.7999992370605}, {"数值"=timestamp(3724657376.000003 s since 1904-01-01), "数值 2"=-38.7999992370605}, {"数值"=timestamp(3724657476.000003 s since 1904-01-01), "数值 2"=-40.5}, {"数值"=timestamp(3724657576.000003 s since 1904-01-01), "数值 2"=-41.0999984741211}, {"数值"=timestamp(3724657676.000003 s since 1904-01-01), "数值 2"=-40.7999992370605}, {"数值"=timestamp(3724657776.000003 s since 1904-01-01), "数值 2"=-39.0}, {"数值"=timestamp(3724657876.000003 s since 1904-01-01), "数值 2"=-38.7000007629395}, {"数值"=timestamp(3724657976.000003 s since 1904-01-01), "数值 2"=90.0999984741211}, {"数值"=timestamp(3724658076.000003 s since 1904-01-01), "数值 2"=85.4000015258789}, {"数值"=timestamp(3724658176.000003 s since 1904-01-01), "数值 2"=85.0999984741211}, {"数值"=timestamp(3724658276.000003 s since 1904-01-01), "数值 2"=85.0999984741211}, {"数值"=timestamp(3724658376.000003 s since 1904-01-01), "数值 2"=85.0999984741211}, {"数值"=timestamp(3724658476.000003 s since 1904-01-01), "数值 2"=85.0999984741211}, {"数值"=timestamp(3724658576.000003 s since 1904-01-01), "数值 2"=85.0}, {"数值"=timestamp(3724658676.000003 s since 1904-01-01), "数值 2"=85.0}, {"数值"=timestamp(3724658776.000003 s since 1904-01-01), "数值 2"=85.0}, {"数值"=timestamp(3724658876.000003 s since 1904-01-01), "数值 2"=85.0}, {"数值"=timestamp(3724658976.000003 s since 1904-01-01), "数值 2"=85.0999984741211}, {"数值"=timestamp(3724659076.000003 s since 1904-01-01), "数值 2"=84.9000015258789}, {"数值"=timestamp(3724659176.000003 s since 1904-01-01), "数值 2"=84.9000015258789}, {"数值"=timestamp(3724659276.000003 s since 1904-01-01), "数值 2"=85.0}, {"数值"=timestamp(3724659376.000003 s since 1904-01-01), "数值 2"=85.0999984741211}, {"数值"=timestamp(3724659476.000003 s since 1904-01-01), "数值 2"=85.0999984741211}, {"数值"=timestamp(3724659576.000003 s since 1904-01-01), "数值 2"=84.9000015258789}, {"数值"=timestamp(3724659676.000003 s since 1904-01-01), "数值 2"=85.0}, {"数值"=timestamp(3724659776.000003 s since 1904-01-01), "数值 2"=-34.7999992370605}, {"数值"=timestamp(3724659876.000003 s since 1904-01-01), "数值 2"=-42.5}, {"数值"=timestamp(3724659976.000003 s since 1904-01-01), "数值 2"=-41.0}, {"数值"=timestamp(3724660076.000003 s since 1904-01-01), "数值 2"=-39.5}, {"数值"=timestamp(3724660176.000003 s since 1904-01-01), "数值 2"=-38.2999992370605}, {"数值"=timestamp(3724660276.000003 s since 1904-01-01), "数值 2"=-38.9000015258789}, {"数值"=timestamp(3724660376.000003 s since 1904-01-01), "数值 2"=-39.7999992370605}, {"数值"=timestamp(3724660476.000003 s since 1904-01-01), "数值 2"=-40.2999992370605}, {"数值"=timestamp(3724660576.000003 s since 1904-01-01), "数值 2"=-40.5}, {"数值"=timestamp(3724660676.000003 s since 1904-01-01), "数值 2"=-40.5999984741211}, {"数值"=timestamp(3724660776.000003 s since 1904-01-01), "数值 2"=-40.5999984741211}, {"数值"=timestamp(3724660876.000003 s since 1904-01-01), "数值 2"=-39.5999984741211}, {"数值"=timestamp(3724660976.000003 s since 1904-01-01), "数值 2"=-38.7999992370605}, {"数值"=timestamp(3724661076.000003 s since 1904-01-01), "数值 2"=-39.7000007629395}, {"数值"=timestamp(3724661176.000003 s since 1904-01-01), "数值 2"=-40.7000007629395}, {"数值"=timestamp(3724661276.000003 s since 1904-01-01), "数值 2"=-40.7999992370605}, {"数值"=timestamp(3724661376.000003 s since 1904-01-01), "数值 2"=-40.2000007629395}, {"数值"=timestamp(3724661476.000003 s since 1904-01-01), "数值 2"=-38.7999992370605}, {"数值"=timestamp(3724661576.000003 s since 1904-01-01), "数值 2"=-39.5}, {"数值"=timestamp(3724661676.000003 s since 1904-01-01), "数值 2"=-40.7000007629395}, {"数值"=timestamp(3724661776.000003 s since 1904-01-01), "数值 2"=-41.0}, {"数值"=timestamp(3724661876.000003 s since 1904-01-01), "数值 2"=-40.2000007629395}, {"数值"=timestamp(3724661976.000003 s since 1904-01-01), "数值 2"=-38.7999992370605}, {"数值"=timestamp(3724662076.000003 s since 1904-01-01), "数值 2"=-39.2000007629395}, {"数值"=timestamp(3724662176.000003 s since 1904-01-01), "数值 2"=-40.7000007629395}, {"数值"=timestamp(3724662276.000003 s since 1904-01-01), "数值 2"=-41.0999984741211}, {"数值"=timestamp(3724662376.000003 s since 1904-01-01), "数值 2"=-40.5999984741211}, {"数值"=timestamp(3724662476.000003 s since 1904-01-01), "数值 2"=89.8000030517578}, {"数值"=timestamp(3724662576.000003 s since 1904-01-01), "数值 2"=85.0999984741211}, {"数值"=timestamp(3724662676.000003 s since 1904-01-01), "数值 2"=85.0}, {"数值"=timestamp(3724662776.000003 s since 1904-01-01), "数值 2"=85.0}, {"数值"=timestamp(3724662876.000003 s since 1904-01-01), "数值 2"=85.0999984741211}, {"数值"=timestamp(3724662976.000003 s since 1904-01-01), "数值 2"=85.0}, {"数值"=timestamp(3724663076.000003 s since 1904-01-01), "数值 2"=85.0}, {"数值"=timestamp(3724663176.000003 s since 1904-01-01), "数值 2"=85.0}, {"数值"=timestamp(3724663276.000003 s since 1904-01-01), "数值 2"=85.0}, {"数值"=timestamp(3724663376.000003 s since 1904-01-01), "数值 2"=85.0}, {"数值"=timestamp(3724663476.000003 s since 1904-01-01), "数值 2"=85.0}, {"数值"=timestamp(3724663576.000003 s since 1904-01-01), "数值 2"=85.0}, {"数值"=timestamp(3724663676.000003 s since 1904-01-01), "数值 2"=85.0}, {"数值"=timestamp(3724663776.000003 s since 1904-01-01), "数值 2"=85.0}, {"数值"=timestamp(3724663876.000003 s since 1904-01-01), "数值 2"=85.0}, {"数值"=timestamp(3724663976.000003 s since 1904-01-01), "数值 2"=85.0}, {"数值"=timestamp(3724664076.000003 s since 1904-01-01), "数值 2"=85.0999984741211}, {"数值"=timestamp(3724664176.000003 s since 1904-01-01), "数值 2"=85.0999984741211}, {"数值"=timestamp(3724664276.000003 s since 1904-01-01), "数值 2"=-39.4000015258789}, {"数值"=timestamp(3724664376.000003 s since 1904-01-01), "数值 2"=-42.4000015258789}, {"数值"=timestamp(3724664476.000003 s since 1904-01-01), "数值 2"=-40.7999992370605}, {"数值"=timestamp(3724664576.000003 s since 1904-01-01), "数值 2"=-39.0}, {"数值"=timestamp(3724664676.000003 s since 1904-01-01), "数值 2"=-38.2000007629395}, {"数值"=timestamp(3724664776.000003 s since 1904-01-01), "数值 2"=-38.9000015258789}, {"数值"=timestamp(3724664876.000003 s since 1904-01-01), "数值 2"=-39.9000015258789}, {"数值"=timestamp(3724664976.000003 s since 1904-01-01), "数值 2"=-40.9000015258789}, {"数值"=timestamp(3724665076.000003 s since 1904-01-01), "数值 2"=-40.9000015258789}, {"数值"=timestamp(3724665176.000003 s since 1904-01-01), "数值 2"=-40.0999984741211}, {"数值"=timestamp(3724665276.000003 s since 1904-01-01), "数值 2"=-38.7000007629395}, {"数值"=timestamp(3724665376.000003 s since 1904-01-01), "数值 2"=-39.5}, {"数值"=timestamp(3724665476.000003 s since 1904-01-01), "数值 2"=-40.7999992370605}, {"数值"=timestamp(3724665576.000003 s since 1904-01-01), "数值 2"=-41.2999992370605}, {"数值"=timestamp(3724665676.000003 s since 1904-01-01), "数值 2"=-40.5}, {"数值"=timestamp(3724665776.000003 s since 1904-01-01), "数值 2"=-39.0999984741211}, {"数值"=timestamp(3724665876.000003 s since 1904-01-01), "数值 2"=-38.5999984741211}, {"数值"=timestamp(3724665976.000003 s since 1904-01-01), "数值 2"=-40.2999992370605}, {"数值"=timestamp(3724666076.000003 s since 1904-01-01), "数值 2"=-41.0}, {"数值"=timestamp(3724666176.000003 s since 1904-01-01), "数值 2"=-41.0}, {"数值"=timestamp(3724666276.000003 s since 1904-01-01), "数值 2"=-40.0999984741211}, {"数值"=timestamp(3724666376.000003 s since 1904-01-01), "数值 2"=-38.5999984741211}, {"数值"=timestamp(3724666476.000003 s since 1904-01-01), "数值 2"=-39.2000007629395}, {"数值"=timestamp(3724666576.000003 s since 1904-01-01), "数值 2"=-40.7000007629395}, {"数值"=timestamp(3724666676.000003 s since 1904-01-01), "数值 2"=-41.0999984741211}, {"数值"=timestamp(3724666776.000003 s since 1904-01-01), "数值 2"=-40.2999992370605}, {"数值"=timestamp(3724666876.000003 s since 1904-01-01), "数值 2"=-38.9000015258789}, {"数值"=timestamp(3724666976.000003 s since 1904-01-01), "数值 2"=88.1999969482422}, {"数值"=timestamp(3724667076.000003 s since 1904-01-01), "数值 2"=85.1999969482422}, {"数值"=timestamp(3724667176.000003 s since 1904-01-01), "数值 2"=85.0999984741211}, {"数值"=timestamp(3724667276.000003 s since 1904-01-01), "数值 2"=85.0999984741211}, {"数值"=timestamp(3724667376.000003 s since 1904-01-01), "数值 2"=84.9000015258789}, {"数值"=timestamp(3724667476.000003 s since 1904-01-01), "数值 2"=85.0}, {"数值"=timestamp(3724667576.000003 s since 1904-01-01), "数值 2"=85.0}, {"数值"=timestamp(3724667676.000003 s since 1904-01-01), "数值 2"=85.0}, {"数值"=timestamp(3724667776.000003 s since 1904-01-01), "数值 2"=85.0}, {"数值"=timestamp(3724667876.000003 s since 1904-01-01), "数值 2"=85.0}, {"数值"=timestamp(3724667976.000003 s since 1904-01-01), "数值 2"=85.0}, {"数值"=timestamp(3724668076.000003 s since 1904-01-01), "数值 2"=85.0}, {"数值"=timestamp(3724668176.000003 s since 1904-01-01), "数值 2"=85.0}, {"数值"=timestamp(3724668276.000003 s since 1904-01-01), "数值 2"=84.9000015258789}, {"数值"=timestamp(3724668376.000003 s since 1904-01-01), "数值 2"=84.9000015258789}, {"数值"=timestamp(3724668476.000003 s since 1904-01-01), "数值 2"=85.0999984741211}, {"数值"=timestamp(3724668576.000003 s since 1904-01-01), "数值 2"=85.0999984741211}, {"数值"=timestamp(3724668676.000003 s since 1904-01-01), "数值 2"=85.0}, {"数值"=timestamp(3724668776.000003 s since 1904-01-01), "数值 2"=-42.0}, {"数值"=timestamp(3724668876.000003 s since 1904-01-01), "数值 2"=-41.4000015258789}, {"数值"=timestamp(3724668976.000003 s since 1904-01-01), "数值 2"=-40.7000007629395}, {"数值"=timestamp(3724669076.000003 s since 1904-01-01), "数值 2"=-39.5999984741211}, {"数值"=timestamp(3724669176.000003 s since 1904-01-01), "数值 2"=-38.0}, {"数值"=timestamp(3724669276.000003 s since 1904-01-01), "数值 2"=-38.5999984741211}, {"数值"=timestamp(3724669376.000003 s since 1904-01-01), "数值 2"=-40.2000007629395}, {"数值"=timestamp(3724669476.000003 s since 1904-01-01), "数值 2"=-41.0}, {"数值"=timestamp(3724669576.000003 s since 1904-01-01), "数值 2"=-41.0999984741211}, {"数值"=timestamp(3724669676.000003 s since 1904-01-01), "数值 2"=-39.7000007629395}, {"数值"=timestamp(3724669776.000003 s since 1904-01-01), "数值 2"=-38.5999984741211}, {"数值"=timestamp(3724669876.000003 s since 1904-01-01), "数值 2"=-39.2999992370605}, {"数值"=timestamp(3724669976.000003 s since 1904-01-01), "数值 2"=-40.7999992370605}, {"数值"=timestamp(3724670076.000003 s since 1904-01-01), "数值 2"=-41.0}, {"数值"=timestamp(3724670176.000003 s since 1904-01-01), "数值 2"=-40.4000015258789}, {"数值"=timestamp(3724670276.000003 s since 1904-01-01), "数值 2"=-38.7000007629395}, {"数值"=timestamp(3724670376.000003 s since 1904-01-01), "数值 2"=-39.0999984741211}, {"数值"=timestamp(3724670476.000003 s since 1904-01-01), "数值 2"=-40.5}, {"数值"=timestamp(3724670576.000003 s since 1904-01-01), "数值 2"=-41.0999984741211}, {"数值"=timestamp(3724670676.000003 s since 1904-01-01), "数值 2"=-40.5}, {"数值"=timestamp(3724670776.000003 s since 1904-01-01), "数值 2"=-39.2999992370605}, {"数值"=timestamp(3724670876.000003 s since 1904-01-01), "数值 2"=-38.7999992370605}, {"数值"=timestamp(3724670976.000003 s since 1904-01-01), "数值 2"=-39.9000015258789}, {"数值"=timestamp(3724671076.000003 s since 1904-01-01), "数值 2"=-40.7999992370605}, {"数值"=timestamp(3724671176.000003 s since 1904-01-01), "数值 2"=-41.0}, {"数值"=timestamp(3724671276.000003 s since 1904-01-01), "数值 2"=-40.2000007629395}, {"数值"=timestamp(3724671376.000003 s since 1904-01-01), "数值 2"=-38.7999992370605}, {"数值"=timestamp(3724671476.000003 s since 1904-01-01), "数值 2"=86.5}, {"数值"=timestamp(3724671576.000003 s since 1904-01-01), "数值 2"=85.1999969482422}, {"数值"=timestamp(3724671676.000003 s since 1904-01-01), "数值 2"=85.0999984741211}, {"数值"=timestamp(3724671776.000003 s since 1904-01-01), "数值 2"=85.0999984741211}, {"数值"=timestamp(3724671876.000003 s since 1904-01-01), "数值 2"=85.0}, {"数值"=timestamp(3724671976.000003 s since 1904-01-01), "数值 2"=85.0}, {"数值"=timestamp(3724672076.000003 s since 1904-01-01), "数值 2"=85.0}, {"数值"=timestamp(3724672176.000003 s since 1904-01-01), "数值 2"=85.0}, {"数值"=timestamp(3724672276.000003 s since 1904-01-01), "数值 2"=85.0}, {"数值"=timestamp(3724672376.000003 s since 1904-01-01), "数值 2"=85.0}, {"数值"=timestamp(3724672476.000003 s since 1904-01-01), "数值 2"=85.0}, {"数值"=timestamp(3724672576.000003 s since 1904-01-01), "数值 2"=85.0}, {"数值"=timestamp(3724672676.000003 s since 1904-01-01), "数值 2"=85.0999984741211}, {"数值"=timestamp(3724672776.000003 s since 1904-01-01), "数值 2"=85.0}, {"数值"=timestamp(3724672876.000003 s since 1904-01-01), "数值 2"=85.0}, {"数值"=timestamp(3724672976.000003 s since 1904-01-01), "数值 2"=84.9000015258789}, {"数值"=timestamp(3724673076.000003 s since 1904-01-01), "数值 2"=85.0}, {"数值"=timestamp(3724673176.000003 s since 1904-01-01), "数值 2"=85.0}, {"数值"=timestamp(3724673276.000003 s since 1904-01-01), "数值 2"=-29.2000007629395}, {"数值"=timestamp(3724673376.000003 s since 1904-01-01), "数值 2"=-41.9000015258789}, {"数值"=timestamp(3724673476.000003 s since 1904-01-01), "数值 2"=-40.9000015258789}, {"数值"=timestamp(3724673576.000003 s since 1904-01-01), "数值 2"=-39.9000015258789}, {"数值"=timestamp(3724673676.000003 s since 1904-01-01), "数值 2"=-38.0999984741211}, {"数值"=timestamp(3724673776.000003 s since 1904-01-01), "数值 2"=-38.7000007629395}, {"数值"=timestamp(3724673876.000003 s since 1904-01-01), "数值 2"=-39.2000007629395}, {"数值"=timestamp(3724673976.000003 s since 1904-01-01), "数值 2"=-40.9000015258789}, {"数值"=timestamp(3724674076.000003 s since 1904-01-01), "数值 2"=-41.0999984741211}, {"数值"=timestamp(3724674176.000003 s since 1904-01-01), "数值 2"=-40.5999984741211}, {"数值"=timestamp(3724674276.000003 s since 1904-01-01), "数值 2"=-38.7000007629395}, {"数值"=timestamp(3724674376.000003 s since 1904-01-01), "数值 2"=-38.9000015258789}, {"数值"=timestamp(3724674476.000003 s since 1904-01-01), "数值 2"=-40.4000015258789}, {"数值"=timestamp(3724674576.000003 s since 1904-01-01), "数值 2"=-41.0}, {"数值"=timestamp(3724674676.000003 s since 1904-01-01), "数值 2"=-40.7000007629395}, {"数值"=timestamp(3724674776.000003 s since 1904-01-01), "数值 2"=-39.2999992370605}, {"数值"=timestamp(3724674876.000003 s since 1904-01-01), "数值 2"=-38.7000007629395}, {"数值"=timestamp(3724674976.000003 s since 1904-01-01), "数值 2"=-40.0999984741211}, {"数值"=timestamp(3724675076.000003 s since 1904-01-01), "数值 2"=-40.9000015258789}, {"数值"=timestamp(3724675176.000003 s since 1904-01-01), "数值 2"=-40.9000015258789}, {"数值"=timestamp(3724675276.000003 s since 1904-01-01), "数值 2"=-40.0}, {"数值"=timestamp(3724675376.000003 s since 1904-01-01), "数值 2"=-38.7000007629395}, {"数值"=timestamp(3724675476.000003 s since 1904-01-01), "数值 2"=-39.4000015258789}, {"数值"=timestamp(3724675576.000003 s since 1904-01-01), "数值 2"=-40.7000007629395}, {"数值"=timestamp(3724675676.000003 s since 1904-01-01), "数值 2"=-41.0}, {"数值"=timestamp(3724675776.000003 s since 1904-01-01), "数值 2"=-40.2999992370605}, {"数值"=timestamp(3724675876.000003 s since 1904-01-01), "数值 2"=-38.7999992370605}, {"数值"=timestamp(3724675976.000003 s since 1904-01-01), "数值 2"=90.5999984741211}, {"数值"=timestamp(3724676076.000003 s since 1904-01-01), "数值 2"=85.1999969482422}, {"数值"=timestamp(3724676176.000003 s since 1904-01-01), "数值 2"=85.0}, {"数值"=timestamp(3724676276.000003 s since 1904-01-01), "数值 2"=85.0}, {"数值"=timestamp(3724676376.000003 s since 1904-01-01), "数值 2"=84.9000015258789}, {"数值"=timestamp(3724676476.000003 s since 1904-01-01), "数值 2"=85.0}, {"数值"=timestamp(3724676576.000003 s since 1904-01-01), "数值 2"=85.0}, {"数值"=timestamp(3724676676.000003 s since 1904-01-01), "数值 2"=85.0}, {"数值"=timestamp(3724676776.000003 s since 1904-01-01), "数值 2"=85.0999984741211}, {"数值"=timestamp(3724676876.000003 s since 1904-01-01), "数值 2"=85.0}, {"数值"=timestamp(3724676976.000003 s since 1904-01-01), "数值 2"=84.9000015258789}, {"数值"=timestamp(3724677076.000003 s since 1904-01-01), "数值 2"=85.0}, {"数值"=timestamp(3724677176.000003 s since 1904-01-01), "数值 2"=85.0}, {"数值"=timestamp(3724677276.000003 s since 1904-01-01), "数值 2"=84.9000015258789}, {"数值"=timestamp(3724677376.000003 s since 1904-01-01), "数值 2"=84.9000015258789}, {"数值"=timestamp(3724677476.000003 s since 1904-01-01), "数值 2"=85.0}, {"数值"=timestamp(3724677576.000003 s since 1904-01-01), "数值 2"=84.9000015258789}, {"数值"=timestamp(3724677676.000003 s since 1904-01-01), "数值 2"=84.9000015258789}, {"数值"=timestamp(3724677776.000003 s since 1904-01-01), "数值 2"=-34.2000007629395}, {"数值"=timestamp(3724677876.000003 s since 1904-01-01), "数值 2"=-41.2999992370605}, {"数值"=timestamp(3724677976.000003 s since 1904-01-01), "数值 2"=-40.7000007629395}, {"数值"=timestamp(3724678076.000003 s since 1904-01-01), "数值 2"=-40.2999992370605}, {"数值"=timestamp(3724678176.000003 s since 1904-01-01), "数值 2"=-38.0}, {"数值"=timestamp(3724678276.000003 s since 1904-01-01), "数值 2"=-38.5}, {"数值"=timestamp(3724678376.000003 s since 1904-01-01), "数值 2"=-39.7999992370605}, {"数值"=timestamp(3724678476.000003 s since 1904-01-01), "数值 2"=-40.7000007629395}, {"数值"=timestamp(3724678576.000003 s since 1904-01-01), "数值 2"=-41.0}, {"数值"=timestamp(3724678676.000003 s since 1904-01-01), "数值 2"=-40.5}, {"数值"=timestamp(3724678776.000003 s since 1904-01-01), "数值 2"=-38.7000007629395}, {"数值"=timestamp(3724678876.000003 s since 1904-01-01), "数值 2"=-39.0}, {"数值"=timestamp(3724678976.000003 s since 1904-01-01), "数值 2"=-40.5}, {"数值"=timestamp(3724679076.000003 s since 1904-01-01), "数值 2"=-41.0999984741211}, {"数值"=timestamp(3724679176.000003 s since 1904-01-01), "数值 2"=-40.7999992370605}, {"数值"=timestamp(3724679276.000003 s since 1904-01-01), "数值 2"=-39.5}, {"数值"=timestamp(3724679376.000003 s since 1904-01-01), "数值 2"=-38.5999984741211}, {"数值"=timestamp(3724679476.000003 s since 1904-01-01), "数值 2"=-40.0}, {"数值"=timestamp(3724679576.000003 s since 1904-01-01), "数值 2"=-41.0}, {"数值"=timestamp(3724679676.000003 s since 1904-01-01), "数值 2"=-40.9000015258789}, {"数值"=timestamp(3724679776.000003 s since 1904-01-01), "数值 2"=-39.9000015258789}, {"数值"=timestamp(3724679876.000003 s since 1904-01-01), "数值 2"=-38.7999992370605}, {"数值"=timestamp(3724679976.000003 s since 1904-01-01), "数值 2"=-39.2999992370605}, {"数值"=timestamp(3724680076.000003 s since 1904-01-01), "数值 2"=-40.7000007629395}, {"数值"=timestamp(3724680176.000003 s since 1904-01-01), "数值 2"=-41.0999984741211}, {"数值"=timestamp(3724680276.000003 s since 1904-01-01), "数值 2"=-40.7000007629395}, {"数值"=timestamp(3724680376.000003 s since 1904-01-01), "数值 2"=-38.9000015258789}, {"数值"=timestamp(3724680476.000003 s since 1904-01-01), "数值 2"=89.9000015258789}, {"数值"=timestamp(3724680576.000003 s since 1904-01-01), "数值 2"=85.1999969482422}, {"数值"=timestamp(3724680676.000003 s since 1904-01-01), "数值 2"=85.0}, {"数值"=timestamp(3724680776.000003 s since 1904-01-01), "数值 2"=85.0}, {"数值"=timestamp(3724680876.000003 s since 1904-01-01), "数值 2"=85.0999984741211}, {"数值"=timestamp(3724680976.000003 s since 1904-01-01), "数值 2"=85.0}, {"数值"=timestamp(3724681076.000003 s since 1904-01-01), "数值 2"=85.0}, {"数值"=timestamp(3724681176.000003 s since 1904-01-01), "数值 2"=85.0}, {"数值"=timestamp(3724681276.000003 s since 1904-01-01), "数值 2"=85.0}, {"数值"=timestamp(3724681376.000003 s since 1904-01-01), "数值 2"=85.0}, {"数值"=timestamp(3724681476.000003 s since 1904-01-01), "数值 2"=85.0}, {"数值"=timestamp(3724681576.000003 s since 1904-01-01), "数值 2"=85.0}, {"数值"=timestamp(3724681676.000003 s since 1904-01-01), "数值 2"=84.9000015258789}, {"数值"=timestamp(3724681776.000003 s since 1904-01-01), "数值 2"=84.9000015258789}, {"数值"=timestamp(3724681876.000003 s since 1904-01-01), "数值 2"=85.0999984741211}, {"数值"=timestamp(3724681976.000003 s since 1904-01-01), "数值 2"=84.9000015258789}, {"数值"=timestamp(3724682076.000003 s since 1904-01-01), "数值 2"=85.0999984741211}, {"数值"=timestamp(3724682176.000003 s since 1904-01-01), "数值 2"=85.0999984741211}, {"数值"=timestamp(3724682276.000003 s since 1904-01-01), "数值 2"=-39.0}, {"数值"=timestamp(3724682376.000003 s since 1904-01-01), "数值 2"=-41.5}, {"数值"=timestamp(3724682476.000003 s since 1904-01-01), "数值 2"=-40.5999984741211}, {"数值"=timestamp(3724682576.000003 s since 1904-01-01), "数值 2"=-39.9000015258789}, {"数值"=timestamp(3724682676.000003 s since 1904-01-01), "数值 2"=-37.9000015258789}, {"数值"=timestamp(3724682776.000003 s since 1904-01-01), "数值 2"=-38.7999992370605}, {"数值"=timestamp(3724682876.000003 s since 1904-01-01), "数值 2"=-39.9000015258789}, {"数值"=timestamp(3724682976.000003 s since 1904-01-01), "数值 2"=-40.9000015258789}, {"数值"=timestamp(3724683076.000003 s since 1904-01-01), "数值 2"=-41.0999984741211}, {"数值"=timestamp(3724683176.000003 s since 1904-01-01), "数值 2"=-40.2999992370605}, {"数值"=timestamp(3724683276.000003 s since 1904-01-01), "数值 2"=-38.9000015258789}, {"数值"=timestamp(3724683376.000003 s since 1904-01-01), "数值 2"=-39.0}, {"数值"=timestamp(3724683476.000003 s since 1904-01-01), "数值 2"=-40.5}, {"数值"=timestamp(3724683576.000003 s since 1904-01-01), "数值 2"=-41.0999984741211}, {"数值"=timestamp(3724683676.000003 s since 1904-01-01), "数值 2"=-40.7000007629395}, {"数值"=timestamp(3724683776.000003 s since 1904-01-01), "数值 2"=-39.5}, {"数值"=timestamp(3724683876.000003 s since 1904-01-01), "数值 2"=-38.5999984741211}, {"数值"=timestamp(3724683976.000003 s since 1904-01-01), "数值 2"=-39.7000007629395}, {"数值"=timestamp(3724684076.000003 s since 1904-01-01), "数值 2"=-40.9000015258789}, {"数值"=timestamp(3724684176.000003 s since 1904-01-01), "数值 2"=-41.0999984741211}, {"数值"=timestamp(3724684276.000003 s since 1904-01-01), "数值 2"=-40.2000007629395}, {"数值"=timestamp(3724684376.000003 s since 1904-01-01), "数值 2"=-38.7999992370605}, {"数值"=timestamp(3724684476.000003 s since 1904-01-01), "数值 2"=-38.7000007629395}, {"数值"=timestamp(3724684576.000003 s since 1904-01-01), "数值 2"=-40.4000015258789}, {"数值"=timestamp(3724684676.000003 s since 1904-01-01), "数值 2"=-41.2000007629395}, {"数值"=timestamp(3724684776.000003 s since 1904-01-01), "数值 2"=-41.0}, {"数值"=timestamp(3724684876.000003 s since 1904-01-01), "数值 2"=-39.7999992370605}, {"数值"=timestamp(3724684976.000003 s since 1904-01-01), "数值 2"=88.5}, {"数值"=timestamp(3724685076.000003 s since 1904-01-01), "数值 2"=85.1999969482422}, {"数值"=timestamp(3724685176.000003 s since 1904-01-01), "数值 2"=85.0}, {"数值"=timestamp(3724685276.000003 s since 1904-01-01), "数值 2"=85.0999984741211}, {"数值"=timestamp(3724685376.000003 s since 1904-01-01), "数值 2"=85.0}, {"数值"=timestamp(3724685476.000003 s since 1904-01-01), "数值 2"=84.9000015258789}, {"数值"=timestamp(3724685576.000003 s since 1904-01-01), "数值 2"=85.0}, {"数值"=timestamp(3724685676.000003 s since 1904-01-01), "数值 2"=85.0}, {"数值"=timestamp(3724685776.000003 s since 1904-01-01), "数值 2"=84.9000015258789}, {"数值"=timestamp(3724685876.000003 s since 1904-01-01), "数值 2"=85.0}, {"数值"=timestamp(3724685976.000003 s since 1904-01-01), "数值 2"=85.0}, {"数值"=timestamp(3724686076.000003 s since 1904-01-01), "数值 2"=85.0999984741211}, {"数值"=timestamp(3724686176.000003 s since 1904-01-01), "数值 2"=85.0}, {"数值"=timestamp(3724686276.000003 s since 1904-01-01), "数值 2"=85.0}, {"数值"=timestamp(3724686376.000003 s since 1904-01-01), "数值 2"=84.9000015258789}, {"数值"=timestamp(3724686476.000003 s since 1904-01-01), "数值 2"=84.9000015258789}, {"数值"=timestamp(3724686576.000003 s since 1904-01-01), "数值 2"=85.0}, {"数值"=timestamp(3724686676.000003 s since 1904-01-01), "数值 2"=85.0}, {"数值"=timestamp(3724686776.000003 s since 1904-01-01), "数值 2"=-41.5}, {"数值"=timestamp(3724686876.000003 s since 1904-01-01), "数值 2"=-41.4000015258789}, {"数值"=timestamp(3724686976.000003 s since 1904-01-01), "数值 2"=-40.5}, {"数值"=timestamp(3724687076.000003 s since 1904-01-01), "数值 2"=-39.7000007629395}, {"数值"=timestamp(3724687176.000003 s since 1904-01-01), "数值 2"=-38.0}, {"数值"=timestamp(3724687276.000003 s since 1904-01-01), "数值 2"=-38.7999992370605}, {"数值"=timestamp(3724687376.000003 s since 1904-01-01), "数值 2"=-39.7999992370605}, {"数值"=timestamp(3724687476.000003 s since 1904-01-01), "数值 2"=-40.9000015258789}, {"数值"=timestamp(3724687576.000003 s since 1904-01-01), "数值 2"=-41.0999984741211}, {"数值"=timestamp(3724687676.000003 s since 1904-01-01), "数值 2"=-40.2999992370605}, {"数值"=timestamp(3724687776.000003 s since 1904-01-01), "数值 2"=-38.9000015258789}, {"数值"=timestamp(3724687876.000003 s since 1904-01-01), "数值 2"=-38.7000007629395}, {"数值"=timestamp(3724687976.000003 s since 1904-01-01), "数值 2"=-40.7000007629395}, {"数值"=timestamp(3724688076.000003 s since 1904-01-01), "数值 2"=-41.0999984741211}, {"数值"=timestamp(3724688176.000003 s since 1904-01-01), "数值 2"=-40.7999992370605}, {"数值"=timestamp(3724688276.000003 s since 1904-01-01), "数值 2"=-39.4000015258789}, {"数值"=timestamp(3724688376.000003 s since 1904-01-01), "数值 2"=-38.5999984741211}, {"数值"=timestamp(3724688476.000003 s since 1904-01-01), "数值 2"=-39.4000015258789}, {"数值"=timestamp(3724688576.000003 s since 1904-01-01), "数值 2"=-40.9000015258789}, {"数值"=timestamp(3724688676.000003 s since 1904-01-01), "数值 2"=-41.0}, {"数值"=timestamp(3724688776.000003 s since 1904-01-01), "数值 2"=-40.4000015258789}, {"数值"=timestamp(3724688876.000003 s since 1904-01-01), "数值 2"=-38.7000007629395}, {"数值"=timestamp(3724688976.000003 s since 1904-01-01), "数值 2"=-39.0}, {"数值"=timestamp(3724689076.000003 s since 1904-01-01), "数值 2"=-40.5}, {"数值"=timestamp(3724689176.000003 s since 1904-01-01), "数值 2"=-41.0999984741211}, {"数值"=timestamp(3724689276.000003 s since 1904-01-01), "数值 2"=-40.7000007629395}, {"数值"=timestamp(3724689376.000003 s since 1904-01-01), "数值 2"=-39.4000015258789}, {"数值"=timestamp(3724689476.000003 s since 1904-01-01), "数值 2"=86.9000015258789}, {"数值"=timestamp(3724689576.000003 s since 1904-01-01), "数值 2"=85.1999969482422}, {"数值"=timestamp(3724689676.000003 s since 1904-01-01), "数值 2"=85.1999969482422}, {"数值"=timestamp(3724689776.000003 s since 1904-01-01), "数值 2"=85.0}, {"数值"=timestamp(3724689876.000003 s since 1904-01-01), "数值 2"=85.0}, {"数值"=timestamp(3724689976.000003 s since 1904-01-01), "数值 2"=85.0}, {"数值"=timestamp(3724690076.000003 s since 1904-01-01), "数值 2"=85.0}, {"数值"=timestamp(3724690176.000003 s since 1904-01-01), "数值 2"=85.0}, {"数值"=timestamp(3724690276.000003 s since 1904-01-01), "数值 2"=85.0}, {"数值"=timestamp(3724690376.000003 s since 1904-01-01), "数值 2"=84.9000015258789}, {"数值"=timestamp(3724690476.000003 s since 1904-01-01), "数值 2"=84.9000015258789}, {"数值"=timestamp(3724690576.000003 s since 1904-01-01), "数值 2"=85.0}, {"数值"=timestamp(3724690676.000003 s since 1904-01-01), "数值 2"=84.9000015258789}, {"数值"=timestamp(3724690776.000003 s since 1904-01-01), "数值 2"=85.0}, {"数值"=timestamp(3724690876.000003 s since 1904-01-01), "数值 2"=85.0}, {"数值"=timestamp(3724690976.000003 s since 1904-01-01), "数值 2"=84.9000015258789}, {"数值"=timestamp(3724691076.000003 s since 1904-01-01), "数值 2"=84.9000015258789}, {"数值"=timestamp(3724691176.000003 s since 1904-01-01), "数值 2"=85.0}, {"数值"=timestamp(3724691276.000003 s since 1904-01-01), "数值 2"=-43.2999992370605}, {"数值"=timestamp(3724691376.000003 s since 1904-01-01), "数值 2"=-41.2999992370605}, {"数值"=timestamp(3724691476.000003 s since 1904-01-01), "数值 2"=-40.5999984741211}, {"数值"=timestamp(3724691576.000003 s since 1904-01-01), "数值 2"=-39.5999984741211}, {"数值"=timestamp(3724691676.000003 s since 1904-01-01), "数值 2"=-38.0999984741211}, {"数值"=timestamp(3724691776.000003 s since 1904-01-01), "数值 2"=-38.7000007629395}, {"数值"=timestamp(3724691876.000003 s since 1904-01-01), "数值 2"=-39.9000015258789}, {"数值"=timestamp(3724691976.000003 s since 1904-01-01), "数值 2"=-41.0}, {"数值"=timestamp(3724692076.000003 s since 1904-01-01), "数值 2"=-41.0999984741211}, {"数值"=timestamp(3724692176.000003 s since 1904-01-01), "数值 2"=-40.0}, {"数值"=timestamp(3724692276.000003 s since 1904-01-01), "数值 2"=-38.7000007629395}, {"数值"=timestamp(3724692376.000003 s since 1904-01-01), "数值 2"=-38.9000015258789}, {"数值"=timestamp(3724692476.000003 s since 1904-01-01), "数值 2"=-40.7000007629395}, {"数值"=timestamp(3724692576.000003 s since 1904-01-01), "数值 2"=-41.0999984741211}, {"数值"=timestamp(3724692676.000003 s since 1904-01-01), "数值 2"=-40.7999992370605}, {"数值"=timestamp(3724692776.000003 s since 1904-01-01), "数值 2"=-39.2000007629395}, {"数值"=timestamp(3724692876.000003 s since 1904-01-01), "数值 2"=-38.7000007629395}, {"数值"=timestamp(3724692976.000003 s since 1904-01-01), "数值 2"=-39.5999984741211}, {"数值"=timestamp(3724693076.000003 s since 1904-01-01), "数值 2"=-41.0}, {"数值"=timestamp(3724693176.000003 s since 1904-01-01), "数值 2"=-41.0}, {"数值"=timestamp(3724693276.000003 s since 1904-01-01), "数值 2"=-40.2999992370605}, {"数值"=timestamp(3724693376.000003 s since 1904-01-01), "数值 2"=-38.5999984741211}, {"数值"=timestamp(3724693476.000003 s since 1904-01-01), "数值 2"=-39.0}, {"数值"=timestamp(3724693576.000003 s since 1904-01-01), "数值 2"=-40.5}, {"数值"=timestamp(3724693676.000003 s since 1904-01-01), "数值 2"=-41.0999984741211}, {"数值"=timestamp(3724693776.000003 s since 1904-01-01), "数值 2"=-40.7000007629395}, {"数值"=timestamp(3724693876.000003 s since 1904-01-01), "数值 2"=-39.4000015258789}, {"数值"=timestamp(3724693976.000003 s since 1904-01-01), "数值 2"=86.1999969482422}, {"数值"=timestamp(3724694076.000003 s since 1904-01-01), "数值 2"=85.1999969482422}, {"数值"=timestamp(3724694176.000003 s since 1904-01-01), "数值 2"=85.1999969482422}, {"数值"=timestamp(3724694276.000003 s since 1904-01-01), "数值 2"=85.0999984741211}, {"数值"=timestamp(3724694376.000003 s since 1904-01-01), "数值 2"=85.0}, {"数值"=timestamp(3724694476.000003 s since 1904-01-01), "数值 2"=85.0}, {"数值"=timestamp(3724694576.000003 s since 1904-01-01), "数值 2"=85.0}, {"数值"=timestamp(3724694676.000003 s since 1904-01-01), "数值 2"=85.0}, {"数值"=timestamp(3724694776.000003 s since 1904-01-01), "数值 2"=84.9000015258789}, {"数值"=timestamp(3724694876.000003 s since 1904-01-01), "数值 2"=85.0}, {"数值"=timestamp(3724694976.000003 s since 1904-01-01), "数值 2"=84.9000015258789}, {"数值"=timestamp(3724695076.000003 s since 1904-01-01), "数值 2"=84.9000015258789}, {"数值"=timestamp(3724695176.000003 s since 1904-01-01), "数值 2"=85.0999984741211}, {"数值"=timestamp(3724695276.000003 s since 1904-01-01), "数值 2"=85.0}, {"数值"=timestamp(3724695376.000003 s since 1904-01-01), "数值 2"=85.0}, {"数值"=timestamp(3724695476.000003 s since 1904-01-01), "数值 2"=85.0999984741211}, {"数值"=timestamp(3724695576.000003 s since 1904-01-01), "数值 2"=84.9000015258789}, {"数值"=timestamp(3724695676.000003 s since 1904-01-01), "数值 2"=85.0}, {"数值"=timestamp(3724695776.000003 s since 1904-01-01), "数值 2"=-33.5999984741211}, {"数值"=timestamp(3724695876.000003 s since 1904-01-01), "数值 2"=-41.7999992370605}, {"数值"=timestamp(3724695976.000003 s since 1904-01-01), "数值 2"=-40.7999992370605}, {"数值"=timestamp(3724696076.000003 s since 1904-01-01), "数值 2"=-39.9000015258789}, {"数值"=timestamp(3724696176.000003 s since 1904-01-01), "数值 2"=-38.2000007629395}, {"数值"=timestamp(3724696276.000003 s since 1904-01-01), "数值 2"=-39.0}, {"数值"=timestamp(3724696376.000003 s since 1904-01-01), "数值 2"=-40.0}, {"数值"=timestamp(3724696476.000003 s since 1904-01-01), "数值 2"=-40.9000015258789}, {"数值"=timestamp(3724696576.000003 s since 1904-01-01), "数值 2"=-40.9000015258789}, {"数值"=timestamp(3724696676.000003 s since 1904-01-01), "数值 2"=-40.0999984741211}, {"数值"=timestamp(3724696776.000003 s since 1904-01-01), "数值 2"=-38.7000007629395}, {"数值"=timestamp(3724696876.000003 s since 1904-01-01), "数值 2"=-39.5999984741211}, {"数值"=timestamp(3724696976.000003 s since 1904-01-01), "数值 2"=-40.5}, {"数值"=timestamp(3724697076.000003 s since 1904-01-01), "数值 2"=-40.9000015258789}, {"数值"=timestamp(3724697176.000003 s since 1904-01-01), "数值 2"=-40.5}, {"数值"=timestamp(3724697276.000003 s since 1904-01-01), "数值 2"=-39.2000007629395}, {"数值"=timestamp(3724697376.000003 s since 1904-01-01), "数值 2"=-38.9000015258789}, {"数值"=timestamp(3724697476.000003 s since 1904-01-01), "数值 2"=-40.4000015258789}, {"数值"=timestamp(3724697576.000003 s since 1904-01-01), "数值 2"=-41.0999984741211}, {"数值"=timestamp(3724697676.000003 s since 1904-01-01), "数值 2"=-40.7999992370605}, {"数值"=timestamp(3724697776.000003 s since 1904-01-01), "数值 2"=-39.5}, {"数值"=timestamp(3724697876.000003 s since 1904-01-01), "数值 2"=-38.5999984741211}, {"数值"=timestamp(3724697976.000003 s since 1904-01-01), "数值 2"=-39.9000015258789}, {"数值"=timestamp(3724698076.000003 s since 1904-01-01), "数值 2"=-40.9000015258789}, {"数值"=timestamp(3724698176.000003 s since 1904-01-01), "数值 2"=-41.0999984741211}, {"数值"=timestamp(3724698276.000003 s since 1904-01-01), "数值 2"=-40.0}, {"数值"=timestamp(3724698376.000003 s since 1904-01-01), "数值 2"=-38.7000007629395}, {"数值"=timestamp(3724698476.000003 s since 1904-01-01), "数值 2"=90.5}, {"数值"=timestamp(3724698576.000003 s since 1904-01-01), "数值 2"=85.3000030517578}, {"数值"=timestamp(3724698676.000003 s since 1904-01-01), "数值 2"=85.0}, {"数值"=timestamp(3724698776.000003 s since 1904-01-01), "数值 2"=85.0}, {"数值"=timestamp(3724698876.000003 s since 1904-01-01), "数值 2"=85.0}, {"数值"=timestamp(3724698976.000003 s since 1904-01-01), "数值 2"=85.0}, {"数值"=timestamp(3724699076.000003 s since 1904-01-01), "数值 2"=85.0}, {"数值"=timestamp(3724699176.000003 s since 1904-01-01), "数值 2"=85.0999984741211}, {"数值"=timestamp(3724699276.000003 s since 1904-01-01), "数值 2"=85.0}, {"数值"=timestamp(3724699376.000003 s since 1904-01-01), "数值 2"=85.0}, {"数值"=timestamp(3724699476.000003 s since 1904-01-01), "数值 2"=85.0999984741211}, {"数值"=timestamp(3724699576.000003 s since 1904-01-01), "数值 2"=85.0999984741211}, {"数值"=timestamp(3724699676.000003 s since 1904-01-01), "数值 2"=84.9000015258789}, {"数值"=timestamp(3724699776.000003 s since 1904-01-01), "数值 2"=85.0}, {"数值"=timestamp(3724699876.000003 s since 1904-01-01), "数值 2"=85.0999984741211}, {"数值"=timestamp(3724699976.000003 s since 1904-01-01), "数值 2"=84.9000015258789}, {"数值"=timestamp(3724700076.000003 s since 1904-01-01), "数值 2"=85.0999984741211}, {"数值"=timestamp(3724700176.000003 s since 1904-01-01), "数值 2"=85.0}, {"数值"=timestamp(3724700276.000003 s since 1904-01-01), "数值 2"=-38.0999984741211}, {"数值"=timestamp(3724700376.000003 s since 1904-01-01), "数值 2"=-41.2000007629395}, {"数值"=timestamp(3724700476.000003 s since 1904-01-01), "数值 2"=-40.7000007629395}, {"数值"=timestamp(3724700576.000003 s since 1904-01-01), "数值 2"=-39.7999992370605}, {"数值"=timestamp(3724700676.000003 s since 1904-01-01), "数值 2"=-38.0999984741211}, {"数值"=timestamp(3724700776.000003 s since 1904-01-01), "数值 2"=-38.7000007629395}, {"数值"=timestamp(3724700876.000003 s since 1904-01-01), "数值 2"=-39.9000015258789}, {"数值"=timestamp(3724700976.000003 s since 1904-01-01), "数值 2"=-41.0}, {"数值"=timestamp(3724701076.000003 s since 1904-01-01), "数值 2"=-41.0}, {"数值"=timestamp(3724701176.000003 s since 1904-01-01), "数值 2"=-40.0999984741211}, {"数值"=timestamp(3724701276.000003 s since 1904-01-01), "数值 2"=-38.5999984741211}, {"数值"=timestamp(3724701376.000003 s since 1904-01-01), "数值 2"=-39.5}, {"数值"=timestamp(3724701476.000003 s since 1904-01-01), "数值 2"=-40.7999992370605}, {"数值"=timestamp(3724701576.000003 s since 1904-01-01), "数值 2"=-41.2000007629395}, {"数值"=timestamp(3724701676.000003 s since 1904-01-01), "数值 2"=-40.2000007629395}, {"数值"=timestamp(3724701776.000003 s since 1904-01-01), "数值 2"=-38.7000007629395}, {"数值"=timestamp(3724701876.000003 s since 1904-01-01), "数值 2"=-38.7999992370605}, {"数值"=timestamp(3724701976.000003 s since 1904-01-01), "数值 2"=-40.5999984741211}, {"数值"=timestamp(3724702076.000003 s since 1904-01-01), "数值 2"=-41.2999992370605}, {"数值"=timestamp(3724702176.000003 s since 1904-01-01), "数值 2"=-40.9000015258789}, {"数值"=timestamp(3724702276.000003 s since 1904-01-01), "数值 2"=-39.2000007629395}, {"数值"=timestamp(3724702376.000003 s since 1904-01-01), "数值 2"=-38.7000007629395}, {"数值"=timestamp(3724702476.000003 s since 1904-01-01), "数值 2"=-39.5}, {"数值"=timestamp(3724702576.000003 s since 1904-01-01), "数值 2"=-41.0}, {"数值"=timestamp(3724702676.000003 s since 1904-01-01), "数值 2"=-41.2000007629395}, {"数值"=timestamp(3724702776.000003 s since 1904-01-01), "数值 2"=-40.5}, {"数值"=timestamp(3724702876.000003 s since 1904-01-01), "数值 2"=-38.5999984741211}, {"数值"=timestamp(3724702976.000003 s since 1904-01-01), "数值 2"=89.0}, {"数值"=timestamp(3724703076.000003 s since 1904-01-01), "数值 2"=85.0999984741211}, {"数值"=timestamp(3724703176.000003 s since 1904-01-01), "数值 2"=85.0999984741211}, {"数值"=timestamp(3724703276.000003 s since 1904-01-01), "数值 2"=85.0}, {"数值"=timestamp(3724703376.000003 s since 1904-01-01), "数值 2"=85.0}, {"数值"=timestamp(3724703476.000003 s since 1904-01-01), "数值 2"=85.0}, {"数值"=timestamp(3724703576.000003 s since 1904-01-01), "数值 2"=85.0}, {"数值"=timestamp(3724703676.000003 s since 1904-01-01), "数值 2"=85.0}, {"数值"=timestamp(3724703776.000003 s since 1904-01-01), "数值 2"=84.9000015258789}, {"数值"=timestamp(3724703876.000003 s since 1904-01-01), "数值 2"=85.0999984741211}, {"数值"=timestamp(3724703976.000003 s since 1904-01-01), "数值 2"=85.0}, {"数值"=timestamp(3724704076.000003 s since 1904-01-01), "数值 2"=85.0}, {"数值"=timestamp(3724704176.000003 s since 1904-01-01), "数值 2"=85.0999984741211}, {"数值"=timestamp(3724704276.000003 s since 1904-01-01), "数值 2"=85.0}, {"数值"=timestamp(3724704376.000003 s since 1904-01-01), "数值 2"=85.0}, {"数值"=timestamp(3724704476.000003 s since 1904-01-01), "数值 2"=84.9000015258789}, {"数值"=timestamp(3724704576.000003 s since 1904-01-01), "数值 2"=85.0}, {"数值"=timestamp(3724704676.000003 s since 1904-01-01), "数值 2"=85.0}, {"数值"=timestamp(3724704776.000003 s since 1904-01-01), "数值 2"=-41.0999984741211}, {"数值"=timestamp(3724704876.000003 s since 1904-01-01), "数值 2"=-41.5}, {"数值"=timestamp(3724704976.000003 s since 1904-01-01), "数值 2"=-40.4000015258789}, {"数值"=timestamp(3724705076.000003 s since 1904-01-01), "数值 2"=-39.2000007629395}, {"数值"=timestamp(3724705176.000003 s since 1904-01-01), "数值 2"=-37.9000015258789}, {"数值"=timestamp(3724705276.000003 s since 1904-01-01), "数值 2"=-38.7000007629395}, {"数值"=timestamp(3724705376.000003 s since 1904-01-01), "数值 2"=-39.9000015258789}, {"数值"=timestamp(3724705476.000003 s since 1904-01-01), "数值 2"=-40.5999984741211}, {"数值"=timestamp(3724705576.000003 s since 1904-01-01), "数值 2"=-40.9000015258789}, {"数值"=timestamp(3724705676.000003 s since 1904-01-01), "数值 2"=-40.5}, {"数值"=timestamp(3724705776.000003 s since 1904-01-01), "数值 2"=-39.0}, {"数值"=timestamp(3724705876.000003 s since 1904-01-01), "数值 2"=-39.2000007629395}, {"数值"=timestamp(3724705976.000003 s since 1904-01-01), "数值 2"=-40.7000007629395}, {"数值"=timestamp(3724706076.000003 s since 1904-01-01), "数值 2"=-41.2000007629395}, {"数值"=timestamp(3724706176.000003 s since 1904-01-01), "数值 2"=-40.5999984741211}, {"数值"=timestamp(3724706276.000003 s since 1904-01-01), "数值 2"=-39.2000007629395}, {"数值"=timestamp(3724706376.000003 s since 1904-01-01), "数值 2"=-38.5999984741211}, {"数值"=timestamp(3724706476.000003 s since 1904-01-01), "数值 2"=-40.0999984741211}, {"数值"=timestamp(3724706576.000003 s since 1904-01-01), "数值 2"=-40.9000015258789}, {"数值"=timestamp(3724706676.000003 s since 1904-01-01), "数值 2"=-41.0}, {"数值"=timestamp(3724706776.000003 s since 1904-01-01), "数值 2"=-39.7000007629395}, {"数值"=timestamp(3724706876.000003 s since 1904-01-01), "数值 2"=-38.5999984741211}, {"数值"=timestamp(3724706976.000003 s since 1904-01-01), "数值 2"=-39.2999992370605}, {"数值"=timestamp(3724707076.000003 s since 1904-01-01), "数值 2"=-40.9000015258789}, {"数值"=timestamp(3724707176.000003 s since 1904-01-01), "数值 2"=-41.0999984741211}, {"数值"=timestamp(3724707276.000003 s since 1904-01-01), "数值 2"=-40.4000015258789}, {"数值"=timestamp(3724707376.000003 s since 1904-01-01), "数值 2"=-38.5999984741211}, {"数值"=timestamp(3724707476.000003 s since 1904-01-01), "数值 2"=86.9000015258789}, {"数值"=timestamp(3724707576.000003 s since 1904-01-01), "数值 2"=85.1999969482422}, {"数值"=timestamp(3724707676.000003 s since 1904-01-01), "数值 2"=85.0}, {"数值"=timestamp(3724707776.000003 s since 1904-01-01), "数值 2"=85.0999984741211}, {"数值"=timestamp(3724707876.000003 s since 1904-01-01), "数值 2"=85.0}, {"数值"=timestamp(3724707976.000003 s since 1904-01-01), "数值 2"=85.0}, {"数值"=timestamp(3724708076.000003 s since 1904-01-01), "数值 2"=85.0}, {"数值"=timestamp(3724708176.000003 s since 1904-01-01), "数值 2"=85.0999984741211}, {"数值"=timestamp(3724708276.000003 s since 1904-01-01), "数值 2"=85.0}, {"数值"=timestamp(3724708376.000003 s since 1904-01-01), "数值 2"=85.0}, {"数值"=timestamp(3724708476.000003 s since 1904-01-01), "数值 2"=85.0}, {"数值"=timestamp(3724708576.000003 s since 1904-01-01), "数值 2"=84.9000015258789}, {"数值"=timestamp(3724708676.000003 s since 1904-01-01), "数值 2"=85.0}, {"数值"=timestamp(3724708776.000003 s since 1904-01-01), "数值 2"=85.0}, {"数值"=timestamp(3724708876.000003 s since 1904-01-01), "数值 2"=85.0}, {"数值"=timestamp(3724708976.000003 s since 1904-01-01), "数值 2"=84.9000015258789}, {"数值"=timestamp(3724709076.000003 s since 1904-01-01), "数值 2"=85.0}, {"数值"=timestamp(3724709176.000003 s since 1904-01-01), "数值 2"=85.0}, {"数值"=timestamp(3724709276.000003 s since 1904-01-01), "数值 2"=-42.9000015258789}, {"数值"=timestamp(3724709376.000003 s since 1904-01-01), "数值 2"=-41.5}, {"数值"=timestamp(3724709476.000003 s since 1904-01-01), "数值 2"=-40.5999984741211}, {"数值"=timestamp(3724709576.000003 s since 1904-01-01), "数值 2"=-39.7000007629395}, {"数值"=timestamp(3724709676.000003 s since 1904-01-01), "数值 2"=-38.0}, {"数值"=timestamp(3724709776.000003 s since 1904-01-01), "数值 2"=-38.4000015258789}, {"数值"=timestamp(3724709876.000003 s since 1904-01-01), "数值 2"=-40.0}, {"数值"=timestamp(3724709976.000003 s since 1904-01-01), "数值 2"=-41.0}, {"数值"=timestamp(3724710076.000003 s since 1904-01-01), "数值 2"=-41.0999984741211}, {"数值"=timestamp(3724710176.000003 s since 1904-01-01), "数值 2"=-39.9000015258789}, {"数值"=timestamp(3724710276.000003 s since 1904-01-01), "数值 2"=-38.5999984741211}, {"数值"=timestamp(3724710376.000003 s since 1904-01-01), "数值 2"=-39.2000007629395}, {"数值"=timestamp(3724710476.000003 s since 1904-01-01), "数值 2"=-40.7999992370605}, {"数值"=timestamp(3724710576.000003 s since 1904-01-01), "数值 2"=-41.0999984741211}, {"数值"=timestamp(3724710676.000003 s since 1904-01-01), "数值 2"=-40.5}, {"数值"=timestamp(3724710776.000003 s since 1904-01-01), "数值 2"=-38.7000007629395}, {"数值"=timestamp(3724710876.000003 s since 1904-01-01), "数值 2"=-38.9000015258789}, {"数值"=timestamp(3724710976.000003 s since 1904-01-01), "数值 2"=-40.5}, {"数值"=timestamp(3724711076.000003 s since 1904-01-01), "数值 2"=-41.2000007629395}, {"数值"=timestamp(3724711176.000003 s since 1904-01-01), "数值 2"=-40.7000007629395}, {"数值"=timestamp(3724711276.000003 s since 1904-01-01), "数值 2"=-39.2999992370605}, {"数值"=timestamp(3724711376.000003 s since 1904-01-01), "数值 2"=-38.7000007629395}, {"数值"=timestamp(3724711476.000003 s since 1904-01-01), "数值 2"=-39.7000007629395}, {"数值"=timestamp(3724711576.000003 s since 1904-01-01), "数值 2"=-40.9000015258789}, {"数值"=timestamp(3724711676.000003 s since 1904-01-01), "数值 2"=-41.0999984741211}, {"数值"=timestamp(3724711776.000003 s since 1904-01-01), "数值 2"=-40.0999984741211}, {"数值"=timestamp(3724711876.000003 s since 1904-01-01), "数值 2"=-38.7000007629395}, {"数值"=timestamp(3724711976.000003 s since 1904-01-01), "数值 2"=85.5}, {"数值"=timestamp(3724712076.000003 s since 1904-01-01), "数值 2"=85.3000030517578}, {"数值"=timestamp(3724712176.000003 s since 1904-01-01), "数值 2"=85.0999984741211}, {"数值"=timestamp(3724712276.000003 s since 1904-01-01), "数值 2"=85.0}, {"数值"=timestamp(3724712376.000003 s since 1904-01-01), "数值 2"=85.0}, {"数值"=timestamp(3724712476.000003 s since 1904-01-01), "数值 2"=85.0}, {"数值"=timestamp(3724712576.000003 s since 1904-01-01), "数值 2"=85.0}, {"数值"=timestamp(3724712676.000003 s since 1904-01-01), "数值 2"=85.0}, {"数值"=timestamp(3724712776.000003 s since 1904-01-01), "数值 2"=85.0}, {"数值"=timestamp(3724712876.000003 s since 1904-01-01), "数值 2"=85.0}, {"数值"=timestamp(3724712976.000003 s since 1904-01-01), "数值 2"=85.0}, {"数值"=timestamp(3724713076.000003 s since 1904-01-01), "数值 2"=84.9000015258789}, {"数值"=timestamp(3724713176.000003 s since 1904-01-01), "数值 2"=85.0}, {"数值"=timestamp(3724713276.000003 s since 1904-01-01), "数值 2"=85.0}, {"数值"=timestamp(3724713376.000003 s since 1904-01-01), "数值 2"=85.0}, {"数值"=timestamp(3724713476.000003 s since 1904-01-01), "数值 2"=85.0999984741211}, {"数值"=timestamp(3724713576.000003 s since 1904-01-01), "数值 2"=85.0999984741211}, {"数值"=timestamp(3724713676.000003 s since 1904-01-01), "数值 2"=84.9000015258789}, {"数值"=timestamp(3724713776.000003 s since 1904-01-01), "数值 2"=-44.0}, {"数值"=timestamp(3724713876.000003 s since 1904-01-01), "数值 2"=-41.4000015258789}, {"数值"=timestamp(3724713976.000003 s since 1904-01-01), "数值 2"=-40.5999984741211}, {"数值"=timestamp(3724714076.000003 s since 1904-01-01), "数值 2"=-39.2000007629395}, {"数值"=timestamp(3724714176.000003 s since 1904-01-01), "数值 2"=-37.9000015258789}, {"数值"=timestamp(3724714276.000003 s since 1904-01-01), "数值 2"=-38.7000007629395}, {"数值"=timestamp(3724714376.000003 s since 1904-01-01), "数值 2"=-40.2000007629395}, {"数值"=timestamp(3724714476.000003 s since 1904-01-01), "数值 2"=-41.0999984741211}, {"数值"=timestamp(3724714576.000003 s since 1904-01-01), "数值 2"=-41.0999984741211}, {"数值"=timestamp(3724714676.000003 s since 1904-01-01), "数值 2"=-39.5999984741211}, {"数值"=timestamp(3724714776.000003 s since 1904-01-01), "数值 2"=-38.5999984741211}, {"数值"=timestamp(3724714876.000003 s since 1904-01-01), "数值 2"=-39.2000007629395}, {"数值"=timestamp(3724714976.000003 s since 1904-01-01), "数值 2"=-40.9000015258789}, {"数值"=timestamp(3724715076.000003 s since 1904-01-01), "数值 2"=-41.0999984741211}, {"数值"=timestamp(3724715176.000003 s since 1904-01-01), "数值 2"=-40.5}, {"数值"=timestamp(3724715276.000003 s since 1904-01-01), "数值 2"=-38.5999984741211}, {"数值"=timestamp(3724715376.000003 s since 1904-01-01), "数值 2"=-38.9000015258789}, {"数值"=timestamp(3724715476.000003 s since 1904-01-01), "数值 2"=-40.4000015258789}, {"数值"=timestamp(3724715576.000003 s since 1904-01-01), "数值 2"=-41.0999984741211}, {"数值"=timestamp(3724715676.000003 s since 1904-01-01), "数值 2"=-40.5999984741211}, {"数值"=timestamp(3724715776.000003 s since 1904-01-01), "数值 2"=-39.2999992370605}, {"数值"=timestamp(3724715876.000003 s since 1904-01-01), "数值 2"=-38.7000007629395}, {"数值"=timestamp(3724715976.000003 s since 1904-01-01), "数值 2"=-40.0}, {"数值"=timestamp(3724716076.000003 s since 1904-01-01), "数值 2"=-41.0}, {"数值"=timestamp(3724716176.000003 s since 1904-01-01), "数值 2"=-41.0999984741211}, {"数值"=timestamp(3724716276.000003 s since 1904-01-01), "数值 2"=-39.7999992370605}, {"数值"=timestamp(3724716376.000003 s since 1904-01-01), "数值 2"=-38.5999984741211}, {"数值"=timestamp(3724716476.000003 s since 1904-01-01), "数值 2"=90.4000015258789}, {"数值"=timestamp(3724716576.000003 s since 1904-01-01), "数值 2"=85.1999969482422}, {"数值"=timestamp(3724716676.000003 s since 1904-01-01), "数值 2"=85.0}, {"数值"=timestamp(3724716776.000003 s since 1904-01-01), "数值 2"=85.0}, {"数值"=timestamp(3724716876.000003 s since 1904-01-01), "数值 2"=85.0999984741211}, {"数值"=timestamp(3724716976.000003 s since 1904-01-01), "数值 2"=85.0}, {"数值"=timestamp(3724717076.000003 s since 1904-01-01), "数值 2"=85.0}, {"数值"=timestamp(3724717176.000003 s since 1904-01-01), "数值 2"=85.0}, {"数值"=timestamp(3724717276.000003 s since 1904-01-01), "数值 2"=85.0}, {"数值"=timestamp(3724717376.000003 s since 1904-01-01), "数值 2"=85.0}, {"数值"=timestamp(3724717476.000003 s since 1904-01-01), "数值 2"=84.9000015258789}, {"数值"=timestamp(3724717576.000003 s since 1904-01-01), "数值 2"=85.0}, {"数值"=timestamp(3724717676.000003 s since 1904-01-01), "数值 2"=85.0}, {"数值"=timestamp(3724717776.000003 s since 1904-01-01), "数值 2"=84.9000015258789}, {"数值"=timestamp(3724717876.000003 s since 1904-01-01), "数值 2"=84.9000015258789}, {"数值"=timestamp(3724717976.000003 s since 1904-01-01), "数值 2"=84.9000015258789}, {"数值"=timestamp(3724718076.000003 s since 1904-01-01), "数值 2"=84.9000015258789}, {"数值"=timestamp(3724718176.000003 s since 1904-01-01), "数值 2"=84.9000015258789}, {"数值"=timestamp(3724718276.000003 s since 1904-01-01), "数值 2"=-37.2999992370605}, {"数值"=timestamp(3724718376.000003 s since 1904-01-01), "数值 2"=-41.4000015258789}, {"数值"=timestamp(3724718476.000003 s since 1904-01-01), "数值 2"=-40.5}, {"数值"=timestamp(3724718576.000003 s since 1904-01-01), "数值 2"=-39.9000015258789}, {"数值"=timestamp(3724718676.000003 s since 1904-01-01), "数值 2"=-38.0}, {"数值"=timestamp(3724718776.000003 s since 1904-01-01), "数值 2"=-38.7999992370605}, {"数值"=timestamp(3724718876.000003 s since 1904-01-01), "数值 2"=-39.7999992370605}, {"数值"=timestamp(3724718976.000003 s since 1904-01-01), "数值 2"=-41.2000007629395}, {"数值"=timestamp(3724719076.000003 s since 1904-01-01), "数值 2"=-41.0999984741211}, {"数值"=timestamp(3724719176.000003 s since 1904-01-01), "数值 2"=-40.0999984741211}, {"数值"=timestamp(3724719276.000003 s since 1904-01-01), "数值 2"=-38.5999984741211}, {"数值"=timestamp(3724719376.000003 s since 1904-01-01), "数值 2"=-39.0999984741211}, {"数值"=timestamp(3724719476.000003 s since 1904-01-01), "数值 2"=-40.7999992370605}, {"数值"=timestamp(3724719576.000003 s since 1904-01-01), "数值 2"=-41.0999984741211}, {"数值"=timestamp(3724719676.000003 s since 1904-01-01), "数值 2"=-40.2999992370605}, {"数值"=timestamp(3724719776.000003 s since 1904-01-01), "数值 2"=-38.7999992370605}, {"数值"=timestamp(3724719876.000003 s since 1904-01-01), "数值 2"=-39.0999984741211}, {"数值"=timestamp(3724719976.000003 s since 1904-01-01), "数值 2"=-40.5999984741211}, {"数值"=timestamp(3724720076.000003 s since 1904-01-01), "数值 2"=-41.0999984741211}, {"数值"=timestamp(3724720176.000003 s since 1904-01-01), "数值 2"=-40.5}, {"数值"=timestamp(3724720276.000003 s since 1904-01-01), "数值 2"=-39.0999984741211}, {"数值"=timestamp(3724720376.000003 s since 1904-01-01), "数值 2"=-38.5999984741211}, {"数值"=timestamp(3724720476.000003 s since 1904-01-01), "数值 2"=-40.4000015258789}, {"数值"=timestamp(3724720576.000003 s since 1904-01-01), "数值 2"=-41.0999984741211}, {"数值"=timestamp(3724720676.000003 s since 1904-01-01), "数值 2"=-40.9000015258789}, {"数值"=timestamp(3724720776.000003 s since 1904-01-01), "数值 2"=-39.2999992370605}, {"数值"=timestamp(3724720876.000003 s since 1904-01-01), "数值 2"=-38.5999984741211}, {"数值"=timestamp(3724720976.000003 s since 1904-01-01), "数值 2"=88.1999969482422}, {"数值"=timestamp(3724721076.000003 s since 1904-01-01), "数值 2"=85.4000015258789}, {"数值"=timestamp(3724721176.000003 s since 1904-01-01), "数值 2"=85.0999984741211}, {"数值"=timestamp(3724721276.000003 s since 1904-01-01), "数值 2"=85.0}, {"数值"=timestamp(3724721376.000003 s since 1904-01-01), "数值 2"=84.9000015258789}, {"数值"=timestamp(3724721476.000003 s since 1904-01-01), "数值 2"=85.0999984741211}, {"数值"=timestamp(3724721576.000003 s since 1904-01-01), "数值 2"=85.0}, {"数值"=timestamp(3724721676.000003 s since 1904-01-01), "数值 2"=85.0}, {"数值"=timestamp(3724721776.000003 s since 1904-01-01), "数值 2"=85.0}, {"数值"=timestamp(3724721876.000003 s since 1904-01-01), "数值 2"=85.0}, {"数值"=timestamp(3724721976.000003 s since 1904-01-01), "数值 2"=85.0}, {"数值"=timestamp(3724722076.000003 s since 1904-01-01), "数值 2"=85.0999984741211}, {"数值"=timestamp(3724722176.000003 s since 1904-01-01), "数值 2"=85.0}, {"数值"=timestamp(3724722276.000003 s since 1904-01-01), "数值 2"=85.0}, {"数值"=timestamp(3724722376.000003 s since 1904-01-01), "数值 2"=85.0}, {"数值"=timestamp(3724722476.000003 s since 1904-01-01), "数值 2"=85.0}, {"数值"=timestamp(3724722576.000003 s since 1904-01-01), "数值 2"=84.9000015258789}, {"数值"=timestamp(3724722676.000003 s since 1904-01-01), "数值 2"=85.0}, {"数值"=timestamp(3724722776.000003 s since 1904-01-01), "数值 2"=-40.7000007629395}, {"数值"=timestamp(3724722876.000003 s since 1904-01-01), "数值 2"=-42.0999984741211}, {"数值"=timestamp(3724722976.000003 s since 1904-01-01), "数值 2"=-40.5999984741211}, {"数值"=timestamp(3724723076.000003 s since 1904-01-01), "数值 2"=-39.0999984741211}, {"数值"=timestamp(3724723176.000003 s since 1904-01-01), "数值 2"=-38.0999984741211}, {"数值"=timestamp(3724723276.000003 s since 1904-01-01), "数值 2"=-38.9000015258789}, {"数值"=timestamp(3724723376.000003 s since 1904-01-01), "数值 2"=-39.7000007629395}, {"数值"=timestamp(3724723476.000003 s since 1904-01-01), "数值 2"=-40.5999984741211}, {"数值"=timestamp(3724723576.000003 s since 1904-01-01), "数值 2"=-40.7999992370605}, {"数值"=timestamp(3724723676.000003 s since 1904-01-01), "数值 2"=-40.5999984741211}, {"数值"=timestamp(3724723776.000003 s since 1904-01-01), "数值 2"=-39.4000015258789}, {"数值"=timestamp(3724723876.000003 s since 1904-01-01), "数值 2"=-39.0}, {"数值"=timestamp(3724723976.000003 s since 1904-01-01), "数值 2"=-40.0}, {"数值"=timestamp(3724724076.000003 s since 1904-01-01), "数值 2"=-40.7000007629395}, {"数值"=timestamp(3724724176.000003 s since 1904-01-01), "数值 2"=-40.9000015258789}, {"数值"=timestamp(3724724276.000003 s since 1904-01-01), "数值 2"=-40.0}, {"数值"=timestamp(3724724376.000003 s since 1904-01-01), "数值 2"=-38.7999992370605}, {"数值"=timestamp(3724724476.000003 s since 1904-01-01), "数值 2"=-39.5}, {"数值"=timestamp(3724724576.000003 s since 1904-01-01), "数值 2"=-40.7999992370605}, {"数值"=timestamp(3724724676.000003 s since 1904-01-01), "数值 2"=-41.2000007629395}, {"数值"=timestamp(3724724776.000003 s since 1904-01-01), "数值 2"=-40.2000007629395}, {"数值"=timestamp(3724724876.000003 s since 1904-01-01), "数值 2"=-38.7000007629395}, {"数值"=timestamp(3724724976.000003 s since 1904-01-01), "数值 2"=-38.7999992370605}, {"数值"=timestamp(3724725076.000003 s since 1904-01-01), "数值 2"=-40.7999992370605}, {"数值"=timestamp(3724725176.000003 s since 1904-01-01), "数值 2"=-41.0999984741211}, {"数值"=timestamp(3724725276.000003 s since 1904-01-01), "数值 2"=-40.7999992370605}, {"数值"=timestamp(3724725376.000003 s since 1904-01-01), "数值 2"=-38.9000015258789}, {"数值"=timestamp(3724725476.000003 s since 1904-01-01), "数值 2"=86.8000030517578}, {"数值"=timestamp(3724725576.000003 s since 1904-01-01), "数值 2"=85.4000015258789}, {"数值"=timestamp(3724725676.000003 s since 1904-01-01), "数值 2"=85.0999984741211}, {"数值"=timestamp(3724725776.000003 s since 1904-01-01), "数值 2"=85.0}, {"数值"=timestamp(3724725876.000003 s since 1904-01-01), "数值 2"=85.0}, {"数值"=timestamp(3724725976.000003 s since 1904-01-01), "数值 2"=85.0}, {"数值"=timestamp(3724726076.000003 s since 1904-01-01), "数值 2"=85.0}, {"数值"=timestamp(3724726176.000003 s since 1904-01-01), "数值 2"=85.0}, {"数值"=timestamp(3724726276.000003 s since 1904-01-01), "数值 2"=85.0}, {"数值"=timestamp(3724726376.000003 s since 1904-01-01), "数值 2"=85.0}, {"数值"=timestamp(3724726476.000003 s since 1904-01-01), "数值 2"=85.0}, {"数值"=timestamp(3724726576.000003 s since 1904-01-01), "数值 2"=85.0999984741211}, {"数值"=timestamp(3724726676.000003 s since 1904-01-01), "数值 2"=85.0999984741211}, {"数值"=timestamp(3724726776.000003 s since 1904-01-01), "数值 2"=85.0}, {"数值"=timestamp(3724726876.000003 s since 1904-01-01), "数值 2"=84.9000015258789}, {"数值"=timestamp(3724726976.000003 s since 1904-01-01), "数值 2"=85.0}, {"数值"=timestamp(3724727076.000003 s since 1904-01-01), "数值 2"=85.0}, {"数值"=timestamp(3724727176.000003 s since 1904-01-01), "数值 2"=85.0}, {"数值"=timestamp(3724727276.000003 s since 1904-01-01), "数值 2"=-43.2000007629395}, {"数值"=timestamp(3724727376.000003 s since 1904-01-01), "数值 2"=-41.5999984741211}, {"数值"=timestamp(3724727476.000003 s since 1904-01-01), "数值 2"=-40.5}, {"数值"=timestamp(3724727576.000003 s since 1904-01-01), "数值 2"=-39.5}, {"数值"=timestamp(3724727676.000003 s since 1904-01-01), "数值 2"=-38.0}, {"数值"=timestamp(3724727776.000003 s since 1904-01-01), "数值 2"=-38.7999992370605}, {"数值"=timestamp(3724727876.000003 s since 1904-01-01), "数值 2"=-39.7999992370605}, {"数值"=timestamp(3724727976.000003 s since 1904-01-01), "数值 2"=-40.7999992370605}, {"数值"=timestamp(3724728076.000003 s since 1904-01-01), "数值 2"=-41.0999984741211}, {"数值"=timestamp(3724728176.000003 s since 1904-01-01), "数值 2"=-40.0999984741211}, {"数值"=timestamp(3724728276.000003 s since 1904-01-01), "数值 2"=-38.7999992370605}, {"数值"=timestamp(3724728376.000003 s since 1904-01-01), "数值 2"=-39.4000015258789}, {"数值"=timestamp(3724728476.000003 s since 1904-01-01), "数值 2"=-40.7000007629395}, {"数值"=timestamp(3724728576.000003 s since 1904-01-01), "数值 2"=-41.2999992370605}, {"数值"=timestamp(3724728676.000003 s since 1904-01-01), "数值 2"=-40.5}, {"数值"=timestamp(3724728776.000003 s since 1904-01-01), "数值 2"=-39.2000007629395}, {"数值"=timestamp(3724728876.000003 s since 1904-01-01), "数值 2"=-38.5}, {"数值"=timestamp(3724728976.000003 s since 1904-01-01), "数值 2"=-39.9000015258789}, {"数值"=timestamp(3724729076.000003 s since 1904-01-01), "数值 2"=-40.7000007629395}, {"数值"=timestamp(3724729176.000003 s since 1904-01-01), "数值 2"=-40.9000015258789}, {"数值"=timestamp(3724729276.000003 s since 1904-01-01), "数值 2"=-40.0}, {"数值"=timestamp(3724729376.000003 s since 1904-01-01), "数值 2"=-38.7000007629395}, {"数值"=timestamp(3724729476.000003 s since 1904-01-01), "数值 2"=-39.2000007629395}, {"数值"=timestamp(3724729576.000003 s since 1904-01-01), "数值 2"=-40.9000015258789}, {"数值"=timestamp(3724729676.000003 s since 1904-01-01), "数值 2"=-41.2000007629395}, {"数值"=timestamp(3724729776.000003 s since 1904-01-01), "数值 2"=-40.5}, {"数值"=timestamp(3724729876.000003 s since 1904-01-01), "数值 2"=-38.5999984741211}, {"数值"=timestamp(3724729976.000003 s since 1904-01-01), "数值 2"=85.8000030517578}, {"数值"=timestamp(3724730076.000003 s since 1904-01-01), "数值 2"=85.1999969482422}, {"数值"=timestamp(3724730176.000003 s since 1904-01-01), "数值 2"=85.0}, {"数值"=timestamp(3724730276.000003 s since 1904-01-01), "数值 2"=85.0}, {"数值"=timestamp(3724730376.000003 s since 1904-01-01), "数值 2"=85.0}, {"数值"=timestamp(3724730476.000003 s since 1904-01-01), "数值 2"=85.0}, {"数值"=timestamp(3724730576.000003 s since 1904-01-01), "数值 2"=85.0}, {"数值"=timestamp(3724730676.000003 s since 1904-01-01), "数值 2"=85.0999984741211}, {"数值"=timestamp(3724730776.000003 s since 1904-01-01), "数值 2"=85.0999984741211}, {"数值"=timestamp(3724730876.000003 s since 1904-01-01), "数值 2"=85.0}, {"数值"=timestamp(3724730976.000003 s since 1904-01-01), "数值 2"=85.0}, {"数值"=timestamp(3724731076.000003 s since 1904-01-01), "数值 2"=84.9000015258789}, {"数值"=timestamp(3724731176.000003 s since 1904-01-01), "数值 2"=85.0}, {"数值"=timestamp(3724731276.000003 s since 1904-01-01), "数值 2"=85.0}, {"数值"=timestamp(3724731376.000003 s since 1904-01-01), "数值 2"=84.9000015258789}, {"数值"=timestamp(3724731476.000003 s since 1904-01-01), "数值 2"=85.0}, {"数值"=timestamp(3724731576.000003 s since 1904-01-01), "数值 2"=85.0}, {"数值"=timestamp(3724731676.000003 s since 1904-01-01), "数值 2"=85.0}, {"数值"=timestamp(3724731776.000003 s since 1904-01-01), "数值 2"=-43.7999992370605}, {"数值"=timestamp(3724731876.000003 s since 1904-01-01), "数值 2"=-41.4000015258789}, {"数值"=timestamp(3724731976.000003 s since 1904-01-01), "数值 2"=-40.4000015258789}, {"数值"=timestamp(3724732076.000003 s since 1904-01-01), "数值 2"=-38.9000015258789}, {"数值"=timestamp(3724732176.000003 s since 1904-01-01), "数值 2"=-38.0}, {"数值"=timestamp(3724732276.000003 s since 1904-01-01), "数值 2"=-38.4000015258789}, {"数值"=timestamp(3724732376.000003 s since 1904-01-01), "数值 2"=-40.0999984741211}, {"数值"=timestamp(3724732476.000003 s since 1904-01-01), "数值 2"=-41.0}, {"数值"=timestamp(3724732576.000003 s since 1904-01-01), "数值 2"=-41.0999984741211}, {"数值"=timestamp(3724732676.000003 s since 1904-01-01), "数值 2"=-39.9000015258789}, {"数值"=timestamp(3724732776.000003 s since 1904-01-01), "数值 2"=-38.5999984741211}, {"数值"=timestamp(3724732876.000003 s since 1904-01-01), "数值 2"=-39.0}, {"数值"=timestamp(3724732976.000003 s since 1904-01-01), "数值 2"=-40.7999992370605}, {"数值"=timestamp(3724733076.000003 s since 1904-01-01), "数值 2"=-41.2999992370605}, {"数值"=timestamp(3724733176.000003 s since 1904-01-01), "数值 2"=-40.7000007629395}, {"数值"=timestamp(3724733276.000003 s since 1904-01-01), "数值 2"=-38.9000015258789}, {"数值"=timestamp(3724733376.000003 s since 1904-01-01), "数值 2"=-38.7000007629395}, {"数值"=timestamp(3724733476.000003 s since 1904-01-01), "数值 2"=-40.0}, {"数值"=timestamp(3724733576.000003 s since 1904-01-01), "数值 2"=-41.0}, {"数值"=timestamp(3724733676.000003 s since 1904-01-01), "数值 2"=-40.9000015258789}, {"数值"=timestamp(3724733776.000003 s since 1904-01-01), "数值 2"=-39.7999992370605}, {"数值"=timestamp(3724733876.000003 s since 1904-01-01), "数值 2"=-38.5999984741211}, {"数值"=timestamp(3724733976.000003 s since 1904-01-01), "数值 2"=-39.7000007629395}, {"数值"=timestamp(3724734076.000003 s since 1904-01-01), "数值 2"=-40.7999992370605}, {"数值"=timestamp(3724734176.000003 s since 1904-01-01), "数值 2"=-41.0}, {"数值"=timestamp(3724734276.000003 s since 1904-01-01), "数值 2"=-40.0999984741211}, {"数值"=timestamp(3724734376.000003 s since 1904-01-01), "数值 2"=-38.7000007629395}, {"数值"=timestamp(3724734476.000003 s since 1904-01-01), "数值 2"=84.9000015258789}, {"数值"=timestamp(3724734576.000003 s since 1904-01-01), "数值 2"=85.5}, {"数值"=timestamp(3724734676.000003 s since 1904-01-01), "数值 2"=85.0999984741211}, {"数值"=timestamp(3724734776.000003 s since 1904-01-01), "数值 2"=85.0}, {"数值"=timestamp(3724734876.000003 s since 1904-01-01), "数值 2"=85.0}, {"数值"=timestamp(3724734976.000003 s since 1904-01-01), "数值 2"=85.0}, {"数值"=timestamp(3724735076.000003 s since 1904-01-01), "数值 2"=85.0}, {"数值"=timestamp(3724735176.000003 s since 1904-01-01), "数值 2"=85.0}, {"数值"=timestamp(3724735276.000003 s since 1904-01-01), "数值 2"=85.0}, {"数值"=timestamp(3724735376.000003 s since 1904-01-01), "数值 2"=85.0}, {"数值"=timestamp(3724735476.000003 s since 1904-01-01), "数值 2"=85.0}, {"数值"=timestamp(3724735576.000003 s since 1904-01-01), "数值 2"=85.0}, {"数值"=timestamp(3724735676.000003 s since 1904-01-01), "数值 2"=85.0999984741211}, {"数值"=timestamp(3724735776.000003 s since 1904-01-01), "数值 2"=85.0}, {"数值"=timestamp(3724735876.000003 s since 1904-01-01), "数值 2"=85.0999984741211}, {"数值"=timestamp(3724735976.000003 s since 1904-01-01), "数值 2"=85.0}, {"数值"=timestamp(3724736076.000003 s since 1904-01-01), "数值 2"=84.9000015258789}, {"数值"=timestamp(3724736176.000003 s since 1904-01-01), "数值 2"=84.9000015258789}, {"数值"=timestamp(3724736276.000003 s since 1904-01-01), "数值 2"=-44.2000007629395}, {"数值"=timestamp(3724736376.000003 s since 1904-01-01), "数值 2"=-41.2999992370605}, {"数值"=timestamp(3724736476.000003 s since 1904-01-01), "数值 2"=-40.5}, {"数值"=timestamp(3724736576.000003 s since 1904-01-01), "数值 2"=-38.5}, {"数值"=timestamp(3724736676.000003 s since 1904-01-01), "数值 2"=-38.0}, {"数值"=timestamp(3724736776.000003 s since 1904-01-01), "数值 2"=-38.7999992370605}, {"数值"=timestamp(3724736876.000003 s since 1904-01-01), "数值 2"=-39.9000015258789}, {"数值"=timestamp(3724736976.000003 s since 1904-01-01), "数值 2"=-40.0999984741211}, {"数值"=timestamp(3724737076.000003 s since 1904-01-01), "数值 2"=-40.2000007629395}, {"数值"=timestamp(3724737176.000003 s since 1904-01-01), "数值 2"=-40.2000007629395}, {"数值"=timestamp(3724737276.000003 s since 1904-01-01), "数值 2"=-40.2999992370605}, {"数值"=timestamp(3724737376.000003 s since 1904-01-01), "数值 2"=-40.2000007629395}, {"数值"=timestamp(3724737476.000003 s since 1904-01-01), "数值 2"=-40.2999992370605}, {"数值"=timestamp(3724737576.000003 s since 1904-01-01), "数值 2"=-40.2000007629395}, {"数值"=timestamp(3724737676.000003 s since 1904-01-01), "数值 2"=-40.0999984741211}, {"数值"=timestamp(3724737776.000003 s since 1904-01-01), "数值 2"=-39.5}, {"数值"=timestamp(3724737876.000003 s since 1904-01-01), "数值 2"=-39.2999992370605}, {"数值"=timestamp(3724737976.000003 s since 1904-01-01), "数值 2"=-39.7000007629395}, {"数值"=timestamp(3724738076.000003 s since 1904-01-01), "数值 2"=-40.0}, {"数值"=timestamp(3724738176.000003 s since 1904-01-01), "数值 2"=-40.0}, {"数值"=timestamp(3724738276.000003 s since 1904-01-01), "数值 2"=-40.2000007629395}, {"数值"=timestamp(3724738376.000003 s since 1904-01-01), "数值 2"=-40.2000007629395}, {"数值"=timestamp(3724738476.000003 s since 1904-01-01), "数值 2"=-40.2999992370605}, {"数值"=timestamp(3724738576.000003 s since 1904-01-01), "数值 2"=-40.2000007629395}, {"数值"=timestamp(3724738676.000003 s since 1904-01-01), "数值 2"=-40.0999984741211}, {"数值"=timestamp(3724738776.000003 s since 1904-01-01), "数值 2"=-40.0}, {"数值"=timestamp(3724738876.000003 s since 1904-01-01), "数值 2"=-40.0}, {"数值"=timestamp(3724738976.000003 s since 1904-01-01), "数值 2"=88.8000030517578}, {"数值"=timestamp(3724739076.000003 s since 1904-01-01), "数值 2"=85.3000030517578}, {"数值"=timestamp(3724739176.000003 s since 1904-01-01), "数值 2"=85.0}, {"数值"=timestamp(3724739276.000003 s since 1904-01-01), "数值 2"=85.0999984741211}, {"数值"=timestamp(3724739376.000003 s since 1904-01-01), "数值 2"=85.0999984741211}, {"数值"=timestamp(3724739476.000003 s since 1904-01-01), "数值 2"=84.9000015258789}, {"数值"=timestamp(3724739576.000003 s since 1904-01-01), "数值 2"=85.0}, {"数值"=timestamp(3724739676.000003 s since 1904-01-01), "数值 2"=85.0}, {"数值"=timestamp(3724739776.000003 s since 1904-01-01), "数值 2"=85.0}, {"数值"=timestamp(3724739876.000003 s since 1904-01-01), "数值 2"=84.9000015258789}, {"数值"=timestamp(3724739976.000003 s since 1904-01-01), "数值 2"=85.0999984741211}, {"数值"=timestamp(3724740076.000003 s since 1904-01-01), "数值 2"=85.0999984741211}, {"数值"=timestamp(3724740176.000003 s since 1904-01-01), "数值 2"=85.0999984741211}, {"数值"=timestamp(3724740276.000003 s since 1904-01-01), "数值 2"=85.0}, {"数值"=timestamp(3724740376.000003 s since 1904-01-01), "数值 2"=85.0}, {"数值"=timestamp(3724740476.000003 s since 1904-01-01), "数值 2"=85.0999984741211}, {"数值"=timestamp(3724740576.000003 s since 1904-01-01), "数值 2"=85.0}, {"数值"=timestamp(3724740676.000003 s since 1904-01-01), "数值 2"=85.0999984741211}, {"数值"=timestamp(3724740776.000003 s since 1904-01-01), "数值 2"=-41.0}, {"数值"=timestamp(3724740876.000003 s since 1904-01-01), "数值 2"=-41.7000007629395}, {"数值"=timestamp(3724740976.000003 s since 1904-01-01), "数值 2"=-40.7999992370605}, {"数值"=timestamp(3724741076.000003 s since 1904-01-01), "数值 2"=-40.0}, {"数值"=timestamp(3724741176.000003 s since 1904-01-01), "数值 2"=-38.0999984741211}, {"数值"=timestamp(3724741276.000003 s since 1904-01-01), "数值 2"=-39.2000007629395}, {"数值"=timestamp(3724741376.000003 s since 1904-01-01), "数值 2"=-40.0999984741211}, {"数值"=timestamp(3724741476.000003 s since 1904-01-01), "数值 2"=-41.0}, {"数值"=timestamp(3724741576.000003 s since 1904-01-01), "数值 2"=-40.9000015258789}, {"数值"=timestamp(3724741676.000003 s since 1904-01-01), "数值 2"=-39.7999992370605}, {"数值"=timestamp(3724741776.000003 s since 1904-01-01), "数值 2"=-38.7999992370605}, {"数值"=timestamp(3724741876.000003 s since 1904-01-01), "数值 2"=-39.5}, {"数值"=timestamp(3724741976.000003 s since 1904-01-01), "数值 2"=-40.7999992370605}, {"数值"=timestamp(3724742076.000003 s since 1904-01-01), "数值 2"=-41.0999984741211}, {"数值"=timestamp(3724742176.000003 s since 1904-01-01), "数值 2"=-40.4000015258789}, {"数值"=timestamp(3724742276.000003 s since 1904-01-01), "数值 2"=-38.9000015258789}, {"数值"=timestamp(3724742376.000003 s since 1904-01-01), "数值 2"=-38.9000015258789}, {"数值"=timestamp(3724742476.000003 s since 1904-01-01), "数值 2"=-40.2999992370605}, {"数值"=timestamp(3724742576.000003 s since 1904-01-01), "数值 2"=-41.0999984741211}, {"数值"=timestamp(3724742676.000003 s since 1904-01-01), "数值 2"=-40.7999992370605}, {"数值"=timestamp(3724742776.000003 s since 1904-01-01), "数值 2"=-39.5999984741211}, {"数值"=timestamp(3724742876.000003 s since 1904-01-01), "数值 2"=-38.5}, {"数值"=timestamp(3724742976.000003 s since 1904-01-01), "数值 2"=-39.5999984741211}, {"数值"=timestamp(3724743076.000003 s since 1904-01-01), "数值 2"=-40.9000015258789}, {"数值"=timestamp(3724743176.000003 s since 1904-01-01), "数值 2"=-41.0999984741211}, {"数值"=timestamp(3724743276.000003 s since 1904-01-01), "数值 2"=-40.4000015258789}, {"数值"=timestamp(3724743376.000003 s since 1904-01-01), "数值 2"=-39.0}, {"数值"=timestamp(3724743476.000003 s since 1904-01-01), "数值 2"=87.4000015258789}, {"数值"=timestamp(3724743576.000003 s since 1904-01-01), "数值 2"=85.1999969482422}, {"数值"=timestamp(3724743676.000003 s since 1904-01-01), "数值 2"=85.0999984741211}, {"数值"=timestamp(3724743776.000003 s since 1904-01-01), "数值 2"=85.0999984741211}, {"数值"=timestamp(3724743876.000003 s since 1904-01-01), "数值 2"=85.0}, {"数值"=timestamp(3724743976.000003 s since 1904-01-01), "数值 2"=85.0}, {"数值"=timestamp(3724744076.000003 s since 1904-01-01), "数值 2"=85.0}, {"数值"=timestamp(3724744176.000003 s since 1904-01-01), "数值 2"=85.0}, {"数值"=timestamp(3724744276.000003 s since 1904-01-01), "数值 2"=85.0}, {"数值"=timestamp(3724744376.000003 s since 1904-01-01), "数值 2"=84.9000015258789}, {"数值"=timestamp(3724744476.000003 s since 1904-01-01), "数值 2"=85.0}, {"数值"=timestamp(3724744576.000003 s since 1904-01-01), "数值 2"=85.0}, {"数值"=timestamp(3724744676.000003 s since 1904-01-01), "数值 2"=84.9000015258789}, {"数值"=timestamp(3724744776.000003 s since 1904-01-01), "数值 2"=85.0}, {"数值"=timestamp(3724744876.000003 s since 1904-01-01), "数值 2"=84.9000015258789}, {"数值"=timestamp(3724744976.000003 s since 1904-01-01), "数值 2"=85.0}, {"数值"=timestamp(3724745076.000003 s since 1904-01-01), "数值 2"=85.0}, {"数值"=timestamp(3724745176.000003 s since 1904-01-01), "数值 2"=84.9000015258789}, {"数值"=timestamp(3724745276.000003 s since 1904-01-01), "数值 2"=-42.7000007629395}, {"数值"=timestamp(3724745376.000003 s since 1904-01-01), "数值 2"=-42.2000007629395}, {"数值"=timestamp(3724745476.000003 s since 1904-01-01), "数值 2"=-40.7000007629395}, {"数值"=timestamp(3724745576.000003 s since 1904-01-01), "数值 2"=-39.0999984741211}, {"数值"=timestamp(3724745676.000003 s since 1904-01-01), "数值 2"=-38.2000007629395}, {"数值"=timestamp(3724745776.000003 s since 1904-01-01), "数值 2"=-38.9000015258789}, {"数值"=timestamp(3724745876.000003 s since 1904-01-01), "数值 2"=-40.0999984741211}, {"数值"=timestamp(3724745976.000003 s since 1904-01-01), "数值 2"=-40.2999992370605}, {"数值"=timestamp(3724746076.000003 s since 1904-01-01), "数值 2"=-40.4000015258789}, {"数值"=timestamp(3724746176.000003 s since 1904-01-01), "数值 2"=-40.5}, {"数值"=timestamp(3724746276.000003 s since 1904-01-01), "数值 2"=-40.5}, {"数值"=timestamp(3724746376.000003 s since 1904-01-01), "数值 2"=-39.5}, {"数值"=timestamp(3724746476.000003 s since 1904-01-01), "数值 2"=-38.7999992370605}, {"数值"=timestamp(3724746576.000003 s since 1904-01-01), "数值 2"=-40.0}, {"数值"=timestamp(3724746676.000003 s since 1904-01-01), "数值 2"=-41.0}, {"数值"=timestamp(3724746776.000003 s since 1904-01-01), "数值 2"=-41.0}, {"数值"=timestamp(3724746876.000003 s since 1904-01-01), "数值 2"=-40.0999984741211}, {"数值"=timestamp(3724746976.000003 s since 1904-01-01), "数值 2"=-38.5999984741211}, {"数值"=timestamp(3724747076.000003 s since 1904-01-01), "数值 2"=-39.5}, {"数值"=timestamp(3724747176.000003 s since 1904-01-01), "数值 2"=-40.7999992370605}, {"数值"=timestamp(3724747276.000003 s since 1904-01-01), "数值 2"=-41.0999984741211}, {"数值"=timestamp(3724747376.000003 s since 1904-01-01), "数值 2"=-40.2000007629395}, {"数值"=timestamp(3724747476.000003 s since 1904-01-01), "数值 2"=-38.7000007629395}, {"数值"=timestamp(3724747576.000003 s since 1904-01-01), "数值 2"=-39.2000007629395}, {"数值"=timestamp(3724747676.000003 s since 1904-01-01), "数值 2"=-40.7000007629395}, {"数值"=timestamp(3724747776.000003 s since 1904-01-01), "数值 2"=-41.2000007629395}, {"数值"=timestamp(3724747876.000003 s since 1904-01-01), "数值 2"=-40.2999992370605}, {"数值"=timestamp(3724747976.000003 s since 1904-01-01), "数值 2"=-40.0}, {"数值"=timestamp(3724748076.000003 s since 1904-01-01), "数值 2"=-39.0999984741211}, {"数值"=timestamp(3724748176.000003 s since 1904-01-01), "数值 2"=-37.5}, {"数值"=timestamp(3724748276.000003 s since 1904-01-01), "数值 2"=-36.4000015258789}, {"数值"=timestamp(3724748376.000003 s since 1904-01-01), "数值 2"=-35.5}, {"数值"=timestamp(3724748476.000003 s since 1904-01-01), "数值 2"=-34.2999992370605}, {"数值"=timestamp(3724748576.000003 s since 1904-01-01), "数值 2"=-33.5}, {"数值"=timestamp(3724748676.000003 s since 1904-01-01), "数值 2"=-32.7000007629395}, {"数值"=timestamp(3724748776.000003 s since 1904-01-01), "数值 2"=-31.6000003814697}, {"数值"=timestamp(3724748876.000003 s since 1904-01-01), "数值 2"=-31.0}, {"数值"=timestamp(3724748976.000003 s since 1904-01-01), "数值 2"=-30.2000007629395}, {"数值"=timestamp(3724749076.000003 s since 1904-01-01), "数值 2"=-29.2999992370605}, {"数值"=timestamp(3724749176.000003 s since 1904-01-01), "数值 2"=-28.6000003814697}, {"数值"=timestamp(3724749276.000003 s since 1904-01-01), "数值 2"=-28.0}, {"数值"=timestamp(3724749376.000003 s since 1904-01-01), "数值 2"=-27.2999992370605}, {"数值"=timestamp(3724749476.000003 s since 1904-01-01), "数值 2"=-26.7000007629395}, {"数值"=timestamp(3724749576.000003 s since 1904-01-01), "数值 2"=-26.1000003814697}, {"数值"=timestamp(3724749676.000003 s since 1904-01-01), "数值 2"=-25.2999992370605}, {"数值"=timestamp(3724749776.000003 s since 1904-01-01), "数值 2"=-24.7000007629395}, {"数值"=timestamp(3724749876.000003 s since 1904-01-01), "数值 2"=-24.2999992370605}, {"数值"=timestamp(3724749976.000003 s since 1904-01-01), "数值 2"=-23.5}, {"数值"=timestamp(3724750076.000003 s since 1904-01-01), "数值 2"=-23.0}, {"数值"=timestamp(3724750176.000003 s since 1904-01-01), "数值 2"=-22.5}, {"数值"=timestamp(3724750276.000003 s since 1904-01-01), "数值 2"=-21.7999992370605}, {"数值"=timestamp(3724750376.000003 s since 1904-01-01), "数值 2"=-21.2999992370605}, {"数值"=timestamp(3724750476.000003 s since 1904-01-01), "数值 2"=-20.8999996185303}, {"数值"=timestamp(3724750576.000003 s since 1904-01-01), "数值 2"=-20.2999992370605}, {"数值"=timestamp(3724750676.000003 s since 1904-01-01), "数值 2"=-19.7999992370605}, {"数值"=timestamp(3724750776.000003 s since 1904-01-01), "数值 2"=-19.3999996185303}, {"数值"=timestamp(3724750876.000003 s since 1904-01-01), "数值 2"=-18.7999992370605}, {"数值"=timestamp(3724750976.000003 s since 1904-01-01), "数值 2"=-18.2999992370605}, {"数值"=timestamp(3724751076.000003 s since 1904-01-01), "数值 2"=-17.8999996185303}, {"数值"=timestamp(3724751176.000003 s since 1904-01-01), "数值 2"=-17.3999996185303}, {"数值"=timestamp(3724751276.000003 s since 1904-01-01), "数值 2"=-17.0}, {"数值"=timestamp(3724751376.000003 s since 1904-01-01), "数值 2"=-16.6000003814697}, {"数值"=timestamp(3724751476.000003 s since 1904-01-01), "数值 2"=-16.2000007629395}, {"数值"=timestamp(3724751576.000003 s since 1904-01-01), "数值 2"=-15.6999998092651}, {"数值"=timestamp(3724751676.000003 s since 1904-01-01), "数值 2"=-15.3999996185303}, {"数值"=timestamp(3724751776.000003 s since 1904-01-01), "数值 2"=-15.0}, {"数值"=timestamp(3724751876.000003 s since 1904-01-01), "数值 2"=-14.6000003814697}, {"数值"=timestamp(3724751976.000003 s since 1904-01-01), "数值 2"=-14.3000001907349}, {"数值"=timestamp(3724752076.000003 s since 1904-01-01), "数值 2"=-13.8999996185303}, {"数值"=timestamp(3724752176.000003 s since 1904-01-01), "数值 2"=-13.5}, {"数值"=timestamp(3724752276.000003 s since 1904-01-01), "数值 2"=-13.1999998092651}, {"数值"=timestamp(3724752376.000003 s since 1904-01-01), "数值 2"=-12.8999996185303}, {"数值"=timestamp(3724752476.000003 s since 1904-01-01), "数值 2"=-12.5}, {"数值"=timestamp(3724752576.000003 s since 1904-01-01), "数值 2"=-12.1999998092651}, {"数值"=timestamp(3724752676.000003 s since 1904-01-01), "数值 2"=-11.8999996185303}, {"数值"=timestamp(3724752776.000003 s since 1904-01-01), "数值 2"=-11.5}, {"数值"=timestamp(3724752876.000003 s since 1904-01-01), "数值 2"=-11.1999998092651}, {"数值"=timestamp(3724752976.000003 s since 1904-01-01), "数值 2"=-11.0}, {"数值"=timestamp(3724753076.000003 s since 1904-01-01), "数值 2"=-10.6000003814697}, {"数值"=timestamp(3724753176.000003 s since 1904-01-01), "数值 2"=-10.3000001907349}, {"数值"=timestamp(3724753276.000003 s since 1904-01-01), "数值 2"=-10.1000003814697}, {"数值"=timestamp(3724753376.000003 s since 1904-01-01), "数值 2"=-9.69999980926514}, {"数值"=timestamp(3724753476.000003 s since 1904-01-01), "数值 2"=-9.5}, {"数值"=timestamp(3724753576.000003 s since 1904-01-01), "数值 2"=-9.30000019073486}, {"数值"=timestamp(3724753676.000003 s since 1904-01-01), "数值 2"=-9.0}, {"数值"=timestamp(3724753776.000003 s since 1904-01-01), "数值 2"=-8.69999980926514}, {"数值"=timestamp(3724753876.000003 s since 1904-01-01), "数值 2"=-8.5}, {"数值"=timestamp(3724753976.000003 s since 1904-01-01), "数值 2"=-8.19999980926514}, {"数值"=timestamp(3724754076.000003 s since 1904-01-01), "数值 2"=-7.90000009536743}, {"数值"=timestamp(3724754176.000003 s since 1904-01-01), "数值 2"=-7.69999980926514}, {"数值"=timestamp(3724754276.000003 s since 1904-01-01), "数值 2"=-7.40000009536743}, {"数值"=timestamp(3724754376.000003 s since 1904-01-01), "数值 2"=-7.19999980926514}, {"数值"=timestamp(3724754476.000003 s since 1904-01-01), "数值 2"=-7.0}, {"数值"=timestamp(3724754576.000003 s since 1904-01-01), "数值 2"=-6.69999980926514}, {"数值"=timestamp(3724754676.000003 s since 1904-01-01), "数值 2"=-6.59999990463257}, {"数值"=timestamp(3724754776.000003 s since 1904-01-01), "数值 2"=-6.40000009536743}, {"数值"=timestamp(3724754876.000003 s since 1904-01-01), "数值 2"=-6.09999990463257}, {"数值"=timestamp(3724754976.000003 s since 1904-01-01), "数值 2"=-5.90000009536743}, {"数值"=timestamp(3724755076.000003 s since 1904-01-01), "数值 2"=-5.69999980926514}, {"数值"=timestamp(3724755176.000003 s since 1904-01-01), "数值 2"=-5.5}, {"数值"=timestamp(3724755276.000003 s since 1904-01-01), "数值 2"=-5.30000019073486}, {"数值"=timestamp(3724755376.000003 s since 1904-01-01), "数值 2"=-5.09999990463257}, {"数值"=timestamp(3724755476.000003 s since 1904-01-01), "数值 2"=-4.90000009536743}, {"数值"=timestamp(3724755576.000003 s since 1904-01-01), "数值 2"=-4.69999980926514}, {"数值"=timestamp(3724755676.000003 s since 1904-01-01), "数值 2"=-4.59999990463257}, {"数值"=timestamp(3724755776.000003 s since 1904-01-01), "数值 2"=-4.30000019073486}, {"数值"=timestamp(3724755876.000003 s since 1904-01-01), "数值 2"=-4.19999980926514}, {"数值"=timestamp(3724755976.000003 s since 1904-01-01), "数值 2"=-4.0}, {"数值"=timestamp(3724756076.000003 s since 1904-01-01), "数值 2"=-3.79999995231628}, {"数值"=timestamp(3724756176.000003 s since 1904-01-01), "数值 2"=-3.70000004768372}, {"数值"=timestamp(3724756276.000003 s since 1904-01-01), "数值 2"=-3.5}, {"数值"=timestamp(3724756376.000003 s since 1904-01-01), "数值 2"=-3.29999995231628}, {"数值"=timestamp(3724756476.000003 s since 1904-01-01), "数值 2"=-3.20000004768372}, {"数值"=timestamp(3724756576.000003 s since 1904-01-01), "数值 2"=-3.0}, {"数值"=timestamp(3724756676.000003 s since 1904-01-01), "数值 2"=-2.90000009536743}, {"数值"=timestamp(3724756776.000003 s since 1904-01-01), "数值 2"=-2.70000004768372}, {"数值"=timestamp(3724756876.000003 s since 1904-01-01), "数值 2"=-2.59999990463257}, {"数值"=timestamp(3724756976.000003 s since 1904-01-01), "数值 2"=-2.40000009536743}, {"数值"=timestamp(3724757076.000003 s since 1904-01-01), "数值 2"=-2.29999995231628}, {"数值"=timestamp(3724757176.000003 s since 1904-01-01), "数值 2"=-2.09999990463257}, {"数值"=timestamp(3724757276.000003 s since 1904-01-01), "数值 2"=-2.0}, {"数值"=timestamp(3724757376.000003 s since 1904-01-01), "数值 2"=-1.89999997615814}, {"数值"=timestamp(3724757476.000003 s since 1904-01-01), "数值 2"=-1.70000004768372}, {"数值"=timestamp(3724757576.000003 s since 1904-01-01), "数值 2"=-1.60000002384186}, {"数值"=timestamp(3724757676.000003 s since 1904-01-01), "数值 2"=-1.5}, {"数值"=timestamp(3724757776.000003 s since 1904-01-01), "数值 2"=-1.29999995231628}, {"数值"=timestamp(3724757876.000003 s since 1904-01-01), "数值 2"=-1.20000004768372}, {"数值"=timestamp(3724757976.000003 s since 1904-01-01), "数值 2"=-1.10000002384186}, {"数值"=timestamp(3724758076.000003 s since 1904-01-01), "数值 2"=-1.0}, {"数值"=timestamp(3724758176.000003 s since 1904-01-01), "数值 2"=-0.899999976158142}, {"数值"=timestamp(3724758276.000003 s since 1904-01-01), "数值 2"=-0.800000011920929}, {"数值"=timestamp(3724758376.000003 s since 1904-01-01), "数值 2"=-0.699999988079071}, {"数值"=timestamp(3724758476.000003 s since 1904-01-01), "数值 2"=-0.600000023841858}, {"数值"=timestamp(3724758576.000003 s since 1904-01-01), "数值 2"=-0.5}, {"数值"=timestamp(3724758676.000003 s since 1904-01-01), "数值 2"=-0.400000005960464}, {"数值"=timestamp(3724758776.000003 s since 1904-01-01), "数值 2"=-0.300000011920929}, {"数值"=timestamp(3724758876.000003 s since 1904-01-01), "数值 2"=-0.200000002980232}, {"数值"=timestamp(3724758976.000003 s since 1904-01-01), "数值 2"=-0.100000001490116}, {"数值"=timestamp(3724759076.000003 s since 1904-01-01), "数值 2"=0.0}, {"数值"=timestamp(3724759176.000003 s since 1904-01-01), "数值 2"=0.100000001490116}, {"数值"=timestamp(3724759276.000003 s since 1904-01-01), "数值 2"=0.200000002980232}, {"数值"=timestamp(3724759376.000003 s since 1904-01-01), "数值 2"=0.300000011920929}, {"数值"=timestamp(3724759476.000003 s since 1904-01-01), "数值 2"=0.400000005960464}, {"数值"=timestamp(3724759576.000003 s since 1904-01-01), "数值 2"=0.5}, {"数值"=timestamp(3724759676.000003 s since 1904-01-01), "数值 2"=0.600000023841858}, {"数值"=timestamp(3724759776.000003 s since 1904-01-01), "数值 2"=0.699999988079071}, {"数值"=timestamp(3724759876.000003 s since 1904-01-01), "数值 2"=0.800000011920929}, {"数值"=timestamp(3724759976.000003 s since 1904-01-01), "数值 2"=0.899999976158142}, {"数值"=timestamp(3724760076.000003 s since 1904-01-01), "数值 2"=1.0}, {"数值"=timestamp(3724760176.000003 s since 1904-01-01), "数值 2"=1.10000002384186}, {"数值"=timestamp(3724760276.000003 s since 1904-01-01), "数值 2"=1.20000004768372}, {"数值"=timestamp(3724760376.000003 s since 1904-01-01), "数值 2"=1.29999995231628}, {"数值"=timestamp(3724760476.000003 s since 1904-01-01), "数值 2"=1.39999997615814}, {"数值"=timestamp(3724760576.000003 s since 1904-01-01), "数值 2"=1.39999997615814}, {"数值"=timestamp(3724760676.000003 s since 1904-01-01), "数值 2"=1.5}, {"数值"=timestamp(3724760776.000003 s since 1904-01-01), "数值 2"=1.60000002384186}, {"数值"=timestamp(3724760876.000003 s since 1904-01-01), "数值 2"=1.70000004768372}, {"数值"=timestamp(3724760976.000003 s since 1904-01-01), "数值 2"=1.79999995231628}, {"数值"=timestamp(3724761076.000003 s since 1904-01-01), "数值 2"=1.89999997615814}, {"数值"=timestamp(3724761176.000003 s since 1904-01-01), "数值 2"=1.89999997615814}, {"数值"=timestamp(3724761276.000003 s since 1904-01-01), "数值 2"=2.09999990463257}, {"数值"=timestamp(3724761376.000003 s since 1904-01-01), "数值 2"=2.09999990463257}, {"数值"=timestamp(3724761476.000003 s since 1904-01-01), "数值 2"=2.20000004768372}, {"数值"=timestamp(3724761576.000003 s since 1904-01-01), "数值 2"=2.29999995231628}, {"数值"=timestamp(3724761676.000003 s since 1904-01-01), "数值 2"=2.40000009536743}, {"数值"=timestamp(3724761776.000003 s since 1904-01-01), "数值 2"=2.5}, {"数值"=timestamp(3724761876.000003 s since 1904-01-01), "数值 2"=2.59999990463257}, {"数值"=timestamp(3724761976.000003 s since 1904-01-01), "数值 2"=2.59999990463257}, {"数值"=timestamp(3724762076.000003 s since 1904-01-01), "数值 2"=2.70000004768372}, {"数值"=timestamp(3724762176.000003 s since 1904-01-01), "数值 2"=2.79999995231628}, {"数值"=timestamp(3724762276.000003 s since 1904-01-01), "数值 2"=2.90000009536743}, {"数值"=timestamp(3724762376.000003 s since 1904-01-01), "数值 2"=2.90000009536743}, {"数值"=timestamp(3724762476.000003 s since 1904-01-01), "数值 2"=3.0}, {"数值"=timestamp(3724762576.000003 s since 1904-01-01), "数值 2"=3.09999990463257}, {"数值"=timestamp(3724762676.000003 s since 1904-01-01), "数值 2"=3.20000004768372}, {"数值"=timestamp(3724762776.000003 s since 1904-01-01), "数值 2"=3.29999995231628}, {"数值"=timestamp(3724762876.000003 s since 1904-01-01), "数值 2"=3.29999995231628}, {"数值"=timestamp(3724762976.000003 s since 1904-01-01), "数值 2"=3.40000009536743}, {"数值"=timestamp(3724763076.000003 s since 1904-01-01), "数值 2"=3.5}, {"数值"=timestamp(3724763176.000003 s since 1904-01-01), "数值 2"=3.59999990463257}, {"数值"=timestamp(3724763276.000003 s since 1904-01-01), "数值 2"=3.59999990463257}, {"数值"=timestamp(3724763376.000003 s since 1904-01-01), "数值 2"=3.70000004768372}, {"数值"=timestamp(3724763476.000003 s since 1904-01-01), "数值 2"=3.79999995231628}, {"数值"=timestamp(3724763576.000003 s since 1904-01-01), "数值 2"=3.90000009536743}, {"数值"=timestamp(3724763676.000003 s since 1904-01-01), "数值 2"=4.0}, {"数值"=timestamp(3724763776.000003 s since 1904-01-01), "数值 2"=4.0}, {"数值"=timestamp(3724763876.000003 s since 1904-01-01), "数值 2"=4.09999990463257}, {"数值"=timestamp(3724763976.000003 s since 1904-01-01), "数值 2"=4.19999980926514}, {"数值"=timestamp(3724764076.000003 s since 1904-01-01), "数值 2"=4.30000019073486}, {"数值"=timestamp(3724764176.000003 s since 1904-01-01), "数值 2"=4.30000019073486}, {"数值"=timestamp(3724764276.000003 s since 1904-01-01), "数值 2"=4.40000009536743}, {"数值"=timestamp(3724764376.000003 s since 1904-01-01), "数值 2"=4.5}, {"数值"=timestamp(3724764476.000003 s since 1904-01-01), "数值 2"=4.5}, {"数值"=timestamp(3724764576.000003 s since 1904-01-01), "数值 2"=4.59999990463257}, {"数值"=timestamp(3724764676.000003 s since 1904-01-01), "数值 2"=4.69999980926514}, {"数值"=timestamp(3724764776.000003 s since 1904-01-01), "数值 2"=4.69999980926514}, {"数值"=timestamp(3724764876.000003 s since 1904-01-01), "数值 2"=4.80000019073486}, {"数值"=timestamp(3724764976.000003 s since 1904-01-01), "数值 2"=4.90000009536743}, {"数值"=timestamp(3724765076.000003 s since 1904-01-01), "数值 2"=5.0}, {"数值"=timestamp(3724765176.000003 s since 1904-01-01), "数值 2"=5.0}, {"数值"=timestamp(3724765276.000003 s since 1904-01-01), "数值 2"=5.09999990463257}, {"数值"=timestamp(3724765376.000003 s since 1904-01-01), "数值 2"=5.19999980926514}, {"数值"=timestamp(3724765476.000003 s since 1904-01-01), "数值 2"=5.19999980926514}, {"数值"=timestamp(3724765576.000003 s since 1904-01-01), "数值 2"=5.30000019073486}, {"数值"=timestamp(3724765676.000003 s since 1904-01-01), "数值 2"=5.40000009536743}, {"数值"=timestamp(3724765776.000003 s since 1904-01-01), "数值 2"=5.40000009536743}, {"数值"=timestamp(3724765876.000003 s since 1904-01-01), "数值 2"=5.5}, {"数值"=timestamp(3724765976.000003 s since 1904-01-01), "数值 2"=5.5}, {"数值"=timestamp(3724766076.000003 s since 1904-01-01), "数值 2"=5.59999990463257}, {"数值"=timestamp(3724766176.000003 s since 1904-01-01), "数值 2"=5.69999980926514}, {"数值"=timestamp(3724766276.000003 s since 1904-01-01), "数值 2"=5.69999980926514}, {"数值"=timestamp(3724766376.000003 s since 1904-01-01), "数值 2"=5.80000019073486}, {"数值"=timestamp(3724766476.000003 s since 1904-01-01), "数值 2"=5.90000009536743}, {"数值"=timestamp(3724766576.000003 s since 1904-01-01), "数值 2"=5.90000009536743}, {"数值"=timestamp(3724766676.000003 s since 1904-01-01), "数值 2"=6.0}, {"数值"=timestamp(3724766776.000003 s since 1904-01-01), "数值 2"=6.0}, {"数值"=timestamp(3724766876.000003 s since 1904-01-01), "数值 2"=6.09999990463257}, {"数值"=timestamp(3724766976.000003 s since 1904-01-01), "数值 2"=6.09999990463257}, {"数值"=timestamp(3724767076.000003 s since 1904-01-01), "数值 2"=6.19999980926514}, {"数值"=timestamp(3724767176.000003 s since 1904-01-01), "数值 2"=6.30000019073486}, {"数值"=timestamp(3724767276.000003 s since 1904-01-01), "数值 2"=6.30000019073486}, {"数值"=timestamp(3724767376.000003 s since 1904-01-01), "数值 2"=6.40000009536743}, {"数值"=timestamp(3724767476.000003 s since 1904-01-01), "数值 2"=6.40000009536743}, {"数值"=timestamp(3724767576.000003 s since 1904-01-01), "数值 2"=6.5}, {"数值"=timestamp(3724767676.000003 s since 1904-01-01), "数值 2"=6.5}, {"数值"=timestamp(3724767776.000003 s since 1904-01-01), "数值 2"=6.59999990463257}, {"数值"=timestamp(3724767876.000003 s since 1904-01-01), "数值 2"=6.59999990463257}, {"数值"=timestamp(3724767976.000003 s since 1904-01-01), "数值 2"=6.69999980926514}, {"数值"=timestamp(3724768076.000003 s since 1904-01-01), "数值 2"=6.69999980926514}, {"数值"=timestamp(3724768176.000003 s since 1904-01-01), "数值 2"=6.80000019073486}, {"数值"=timestamp(3724768276.000003 s since 1904-01-01), "数值 2"=6.80000019073486}, {"数值"=timestamp(3724768376.000003 s since 1904-01-01), "数值 2"=6.90000009536743}, {"数值"=timestamp(3724768476.000003 s since 1904-01-01), "数值 2"=6.90000009536743}, {"数值"=timestamp(3724768576.000003 s since 1904-01-01), "数值 2"=7.0}, {"数值"=timestamp(3724768676.000003 s since 1904-01-01), "数值 2"=7.0}, {"数值"=timestamp(3724768776.000003 s since 1904-01-01), "数值 2"=7.09999990463257}, {"数值"=timestamp(3724768876.000003 s since 1904-01-01), "数值 2"=7.09999990463257}, {"数值"=timestamp(3724768976.000003 s since 1904-01-01), "数值 2"=7.19999980926514}, {"数值"=timestamp(3724769076.000003 s since 1904-01-01), "数值 2"=7.19999980926514}, {"数值"=timestamp(3724769176.000003 s since 1904-01-01), "数值 2"=7.30000019073486}, {"数值"=timestamp(3724769276.000003 s since 1904-01-01), "数值 2"=7.30000019073486}, {"数值"=timestamp(3724769376.000003 s since 1904-01-01), "数值 2"=7.40000009536743}, {"数值"=timestamp(3724769476.000003 s since 1904-01-01), "数值 2"=7.40000009536743}, {"数值"=timestamp(3724769576.000003 s since 1904-01-01), "数值 2"=7.5}, {"数值"=timestamp(3724769676.000003 s since 1904-01-01), "数值 2"=7.5}, {"数值"=timestamp(3724769776.000003 s since 1904-01-01), "数值 2"=7.5}, {"数值"=timestamp(3724769876.000003 s since 1904-01-01), "数值 2"=7.59999990463257}, {"数值"=timestamp(3724769976.000003 s since 1904-01-01), "数值 2"=7.59999990463257}, {"数值"=timestamp(3724770076.000003 s since 1904-01-01), "数值 2"=7.69999980926514}, {"数值"=timestamp(3724770176.000003 s since 1904-01-01), "数值 2"=7.69999980926514}, {"数值"=timestamp(3724770276.000003 s since 1904-01-01), "数值 2"=7.80000019073486}, {"数值"=timestamp(3724770376.000003 s since 1904-01-01), "数值 2"=7.80000019073486}, {"数值"=timestamp(3724770476.000003 s since 1904-01-01), "数值 2"=7.90000009536743}, {"数值"=timestamp(3724770576.000003 s since 1904-01-01), "数值 2"=7.90000009536743}, {"数值"=timestamp(3724770676.000003 s since 1904-01-01), "数值 2"=7.90000009536743}, {"数值"=timestamp(3724770776.000003 s since 1904-01-01), "数值 2"=8.0}, {"数值"=timestamp(3724770876.000003 s since 1904-01-01), "数值 2"=8.0}, {"数值"=timestamp(3724770976.000003 s since 1904-01-01), "数值 2"=8.10000038146973}, {"数值"=timestamp(3724771076.000003 s since 1904-01-01), "数值 2"=8.10000038146973}, {"数值"=timestamp(3724771176.000003 s since 1904-01-01), "数值 2"=8.10000038146973}, {"数值"=timestamp(3724771276.000003 s since 1904-01-01), "数值 2"=8.19999980926514}, {"数值"=timestamp(3724771376.000003 s since 1904-01-01), "数值 2"=8.19999980926514}, {"数值"=timestamp(3724771476.000003 s since 1904-01-01), "数值 2"=8.30000019073486}, {"数值"=timestamp(3724771576.000003 s since 1904-01-01), "数值 2"=8.30000019073486}, {"数值"=timestamp(3724771676.000003 s since 1904-01-01), "数值 2"=8.30000019073486}, {"数值"=timestamp(3724771776.000003 s since 1904-01-01), "数值 2"=8.39999961853027}, {"数值"=timestamp(3724771876.000003 s since 1904-01-01), "数值 2"=8.39999961853027}, {"数值"=timestamp(3724771976.000003 s since 1904-01-01), "数值 2"=8.39999961853027}, {"数值"=timestamp(3724772076.000003 s since 1904-01-01), "数值 2"=8.5}, {"数值"=timestamp(3724772176.000003 s since 1904-01-01), "数值 2"=8.5}, {"数值"=timestamp(3724772276.000003 s since 1904-01-01), "数值 2"=8.60000038146973}, {"数值"=timestamp(3724772376.000003 s since 1904-01-01), "数值 2"=8.60000038146973}, {"数值"=timestamp(3724772476.000003 s since 1904-01-01), "数值 2"=8.60000038146973}, {"数值"=timestamp(3724772576.000003 s since 1904-01-01), "数值 2"=8.69999980926514}, {"数值"=timestamp(3724772676.000003 s since 1904-01-01), "数值 2"=8.69999980926514}, {"数值"=timestamp(3724772776.000003 s since 1904-01-01), "数值 2"=8.69999980926514}, {"数值"=timestamp(3724772876.000003 s since 1904-01-01), "数值 2"=8.80000019073486}, {"数值"=timestamp(3724772976.000003 s since 1904-01-01), "数值 2"=8.80000019073486}, {"数值"=timestamp(3724773076.000003 s since 1904-01-01), "数值 2"=8.80000019073486}, {"数值"=timestamp(3724773176.000003 s since 1904-01-01), "数值 2"=8.89999961853027}, {"数值"=timestamp(3724773276.000003 s since 1904-01-01), "数值 2"=8.89999961853027}, {"数值"=timestamp(3724773376.000003 s since 1904-01-01), "数值 2"=8.89999961853027}, {"数值"=timestamp(3724773476.000003 s since 1904-01-01), "数值 2"=9.0}, {"数值"=timestamp(3724773576.000003 s since 1904-01-01), "数值 2"=9.0}, {"数值"=timestamp(3724773676.000003 s since 1904-01-01), "数值 2"=9.0}, {"数值"=timestamp(3724773776.000003 s since 1904-01-01), "数值 2"=9.10000038146973}, {"数值"=timestamp(3724773876.000003 s since 1904-01-01), "数值 2"=9.10000038146973}, {"数值"=timestamp(3724773976.000003 s since 1904-01-01), "数值 2"=9.10000038146973}, {"数值"=timestamp(3724774076.000003 s since 1904-01-01), "数值 2"=9.19999980926514}, {"数值"=timestamp(3724774176.000003 s since 1904-01-01), "数值 2"=9.19999980926514}, {"数值"=timestamp(3724774276.000003 s since 1904-01-01), "数值 2"=9.19999980926514}, {"数值"=timestamp(3724774376.000003 s since 1904-01-01), "数值 2"=9.30000019073486}, {"数值"=timestamp(3724774476.000003 s since 1904-01-01), "数值 2"=9.30000019073486}, {"数值"=timestamp(3724774576.000003 s since 1904-01-01), "数值 2"=9.30000019073486}, {"数值"=timestamp(3724774676.000003 s since 1904-01-01), "数值 2"=9.39999961853027}, {"数值"=timestamp(3724774776.000003 s since 1904-01-01), "数值 2"=9.39999961853027}, {"数值"=timestamp(3724774876.000003 s since 1904-01-01), "数值 2"=9.39999961853027}, {"数值"=timestamp(3724774976.000003 s since 1904-01-01), "数值 2"=9.5}, {"数值"=timestamp(3724775076.000003 s since 1904-01-01), "数值 2"=9.5}, {"数值"=timestamp(3724775176.000003 s since 1904-01-01), "数值 2"=9.5}, {"数值"=timestamp(3724775276.000003 s since 1904-01-01), "数值 2"=9.60000038146973}, {"数值"=timestamp(3724775376.000003 s since 1904-01-01), "数值 2"=9.60000038146973}, {"数值"=timestamp(3724775476.000003 s since 1904-01-01), "数值 2"=9.60000038146973}, {"数值"=timestamp(3724775576.000003 s since 1904-01-01), "数值 2"=9.69999980926514}, {"数值"=timestamp(3724775676.000003 s since 1904-01-01), "数值 2"=9.69999980926514}, {"数值"=timestamp(3724775776.000003 s since 1904-01-01), "数值 2"=9.69999980926514}, {"数值"=timestamp(3724775876.000003 s since 1904-01-01), "数值 2"=9.69999980926514}, {"数值"=timestamp(3724775976.000003 s since 1904-01-01), "数值 2"=9.80000019073486}, {"数值"=timestamp(3724776076.000003 s since 1904-01-01), "数值 2"=9.80000019073486}, {"数值"=timestamp(3724776176.000003 s since 1904-01-01), "数值 2"=9.80000019073486}, {"数值"=timestamp(3724776276.000003 s since 1904-01-01), "数值 2"=9.89999961853027}, {"数值"=timestamp(3724776376.000003 s since 1904-01-01), "数值 2"=9.89999961853027}, {"数值"=timestamp(3724776476.000003 s since 1904-01-01), "数值 2"=9.89999961853027}, {"数值"=timestamp(3724776576.000003 s since 1904-01-01), "数值 2"=9.89999961853027}, {"数值"=timestamp(3724776676.000003 s since 1904-01-01), "数值 2"=10.0}, {"数值"=timestamp(3724776776.000003 s since 1904-01-01), "数值 2"=10.0}, {"数值"=timestamp(3724776876.000003 s since 1904-01-01), "数值 2"=10.0}, {"数值"=timestamp(3724776976.000003 s since 1904-01-01), "数值 2"=10.0}, {"数值"=timestamp(3724777076.000003 s since 1904-01-01), "数值 2"=10.1000003814697}, {"数值"=timestamp(3724777176.000003 s since 1904-01-01), "数值 2"=10.1000003814697}, {"数值"=timestamp(3724777276.000003 s since 1904-01-01), "数值 2"=10.1000003814697}, {"数值"=timestamp(3724777376.000003 s since 1904-01-01), "数值 2"=10.1999998092651}, {"数值"=timestamp(3724777476.000003 s since 1904-01-01), "数值 2"=10.1999998092651}, {"数值"=timestamp(3724777576.000003 s since 1904-01-01), "数值 2"=10.1999998092651}, {"数值"=timestamp(3724777676.000003 s since 1904-01-01), "数值 2"=10.1999998092651}, {"数值"=timestamp(3724777776.000003 s since 1904-01-01), "数值 2"=10.3000001907349}, {"数值"=timestamp(3724777876.000003 s since 1904-01-01), "数值 2"=10.3000001907349}, {"数值"=timestamp(3724777976.000003 s since 1904-01-01), "数值 2"=10.3000001907349}, {"数值"=timestamp(3724778076.000003 s since 1904-01-01), "数值 2"=10.3000001907349}, {"数值"=timestamp(3724778176.000003 s since 1904-01-01), "数值 2"=10.3999996185303}, {"数值"=timestamp(3724778276.000003 s since 1904-01-01), "数值 2"=10.3999996185303}, {"数值"=timestamp(3724778376.000003 s since 1904-01-01), "数值 2"=10.3999996185303}, {"数值"=timestamp(3724778476.000003 s since 1904-01-01), "数值 2"=10.3999996185303}, {"数值"=timestamp(3724778576.000003 s since 1904-01-01), "数值 2"=10.5}, {"数值"=timestamp(3724778676.000003 s since 1904-01-01), "数值 2"=10.5}, {"数值"=timestamp(3724778776.000003 s since 1904-01-01), "数值 2"=10.5}, {"数值"=timestamp(3724778876.000003 s since 1904-01-01), "数值 2"=10.5}, {"数值"=timestamp(3724778976.000003 s since 1904-01-01), "数值 2"=10.6000003814697}, {"数值"=timestamp(3724779076.000003 s since 1904-01-01), "数值 2"=10.6000003814697}, {"数值"=timestamp(3724779176.000003 s since 1904-01-01), "数值 2"=10.6000003814697}, {"数值"=timestamp(3724779276.000003 s since 1904-01-01), "数值 2"=10.6000003814697}, {"数值"=timestamp(3724779376.000003 s since 1904-01-01), "数值 2"=10.6999998092651}, {"数值"=timestamp(3724779476.000003 s since 1904-01-01), "数值 2"=10.6999998092651}, {"数值"=timestamp(3724779576.000003 s since 1904-01-01), "数值 2"=10.6999998092651}, {"数值"=timestamp(3724779676.000003 s since 1904-01-01), "数值 2"=10.6999998092651}, {"数值"=timestamp(3724779776.000003 s since 1904-01-01), "数值 2"=10.6999998092651}, {"数值"=timestamp(3724779876.000003 s since 1904-01-01), "数值 2"=10.8000001907349}, {"数值"=timestamp(3724779976.000003 s since 1904-01-01), "数值 2"=10.8000001907349}, {"数值"=timestamp(3724780076.000003 s since 1904-01-01), "数值 2"=10.8000001907349}, {"数值"=timestamp(3724780176.000003 s since 1904-01-01), "数值 2"=10.8000001907349}, {"数值"=timestamp(3724780276.000003 s since 1904-01-01), "数值 2"=10.8999996185303}, {"数值"=timestamp(3724780376.000003 s since 1904-01-01), "数值 2"=10.8999996185303}, {"数值"=timestamp(3724780476.000003 s since 1904-01-01), "数值 2"=10.8999996185303}, {"数值"=timestamp(3724780576.000003 s since 1904-01-01), "数值 2"=10.8999996185303}, {"数值"=timestamp(3724780676.000003 s since 1904-01-01), "数值 2"=10.8999996185303}, {"数值"=timestamp(3724780776.000003 s since 1904-01-01), "数值 2"=11.0}, {"数值"=timestamp(3724780876.000003 s since 1904-01-01), "数值 2"=11.0}, {"数值"=timestamp(3724780976.000003 s since 1904-01-01), "数值 2"=11.0}, {"数值"=timestamp(3724781076.000003 s since 1904-01-01), "数值 2"=11.0}, {"数值"=timestamp(3724781176.000003 s since 1904-01-01), "数值 2"=11.1000003814697}, {"数值"=timestamp(3724781276.000003 s since 1904-01-01), "数值 2"=11.1000003814697}, {"数值"=timestamp(3724781376.000003 s since 1904-01-01), "数值 2"=11.1000003814697}, {"数值"=timestamp(3724781476.000003 s since 1904-01-01), "数值 2"=11.1000003814697}, {"数值"=timestamp(3724781576.000003 s since 1904-01-01), "数值 2"=11.1000003814697}, {"数值"=timestamp(3724781676.000003 s since 1904-01-01), "数值 2"=11.1999998092651}, {"数值"=timestamp(3724781776.000003 s since 1904-01-01), "数值 2"=11.1999998092651}, {"数值"=timestamp(3724781876.000003 s since 1904-01-01), "数值 2"=11.1999998092651}, {"数值"=timestamp(3724781976.000003 s since 1904-01-01), "数值 2"=11.1999998092651}, {"数值"=timestamp(3724782076.000003 s since 1904-01-01), "数值 2"=11.3000001907349}, {"数值"=timestamp(3724782176.000003 s since 1904-01-01), "数值 2"=11.3000001907349}, {"数值"=timestamp(3724782276.000003 s since 1904-01-01), "数值 2"=11.3000001907349}, {"数值"=timestamp(3724782376.000003 s since 1904-01-01), "数值 2"=11.3000001907349}, {"数值"=timestamp(3724782476.000003 s since 1904-01-01), "数值 2"=11.3000001907349}, {"数值"=timestamp(3724782576.000003 s since 1904-01-01), "数值 2"=11.3999996185303}, {"数值"=timestamp(3724782676.000003 s since 1904-01-01), "数值 2"=11.3999996185303}, {"数值"=timestamp(3724782776.000003 s since 1904-01-01), "数值 2"=11.3999996185303}, {"数值"=timestamp(3724782876.000003 s since 1904-01-01), "数值 2"=11.3999996185303}, {"数值"=timestamp(3724782976.000003 s since 1904-01-01), "数值 2"=11.3999996185303}, {"数值"=timestamp(3724783076.000003 s since 1904-01-01), "数值 2"=11.5}, {"数值"=timestamp(3724783176.000003 s since 1904-01-01), "数值 2"=11.5}, {"数值"=timestamp(3724783276.000003 s since 1904-01-01), "数值 2"=11.5}, {"数值"=timestamp(3724783376.000003 s since 1904-01-01), "数值 2"=11.5}, {"数值"=timestamp(3724783476.000003 s since 1904-01-01), "数值 2"=11.5}, {"数值"=timestamp(3724783576.000003 s since 1904-01-01), "数值 2"=11.6000003814697}, {"数值"=timestamp(3724783676.000003 s since 1904-01-01), "数值 2"=11.6000003814697}, {"数值"=timestamp(3724783776.000003 s since 1904-01-01), "数值 2"=11.6000003814697}, {"数值"=timestamp(3724783876.000003 s since 1904-01-01), "数值 2"=11.6000003814697}, {"数值"=timestamp(3724783976.000003 s since 1904-01-01), "数值 2"=11.6000003814697}, {"数值"=timestamp(3724784076.000003 s since 1904-01-01), "数值 2"=11.6999998092651}, {"数值"=timestamp(3724784176.000003 s since 1904-01-01), "数值 2"=11.6999998092651}, {"数值"=timestamp(3724784276.000003 s since 1904-01-01), "数值 2"=11.6999998092651}, {"数值"=timestamp(3724784376.000003 s since 1904-01-01), "数值 2"=11.6999998092651}, {"数值"=timestamp(3724784476.000003 s since 1904-01-01), "数值 2"=11.6999998092651}, {"数值"=timestamp(3724784576.000003 s since 1904-01-01), "数值 2"=11.8000001907349}, {"数值"=timestamp(3724784676.000003 s since 1904-01-01), "数值 2"=11.8000001907349}, {"数值"=timestamp(3724784776.000003 s since 1904-01-01), "数值 2"=11.8000001907349}, {"数值"=timestamp(3724784876.000003 s since 1904-01-01), "数值 2"=11.8000001907349}, {"数值"=timestamp(3724784976.000003 s since 1904-01-01), "数值 2"=11.8000001907349}, {"数值"=timestamp(3724785076.000003 s since 1904-01-01), "数值 2"=11.8999996185303}, {"数值"=timestamp(3724785176.000003 s since 1904-01-01), "数值 2"=11.8999996185303}, {"数值"=timestamp(3724785276.000003 s since 1904-01-01), "数值 2"=11.8999996185303}, {"数值"=timestamp(3724785376.000003 s since 1904-01-01), "数值 2"=11.8999996185303}, {"数值"=timestamp(3724785476.000003 s since 1904-01-01), "数值 2"=11.8999996185303}, {"数值"=timestamp(3724785576.000003 s since 1904-01-01), "数值 2"=11.8999996185303}, {"数值"=timestamp(3724785676.000003 s since 1904-01-01), "数值 2"=12.0}, {"数值"=timestamp(3724785776.000003 s since 1904-01-01), "数值 2"=12.0}, {"数值"=timestamp(3724785876.000003 s since 1904-01-01), "数值 2"=12.0}, {"数值"=timestamp(3724785976.000003 s since 1904-01-01), "数值 2"=12.0}, {"数值"=timestamp(3724786076.000003 s since 1904-01-01), "数值 2"=12.0}, {"数值"=timestamp(3724786176.000003 s since 1904-01-01), "数值 2"=12.1000003814697}, {"数值"=timestamp(3724786276.000003 s since 1904-01-01), "数值 2"=12.1000003814697}, {"数值"=timestamp(3724786376.000003 s since 1904-01-01), "数值 2"=12.1000003814697}, {"数值"=timestamp(3724786476.000003 s since 1904-01-01), "数值 2"=12.1000003814697}, {"数值"=timestamp(3724786576.000003 s since 1904-01-01), "数值 2"=12.1000003814697}, {"数值"=timestamp(3724786676.000003 s since 1904-01-01), "数值 2"=12.1000003814697}, {"数值"=timestamp(3724786776.000003 s since 1904-01-01), "数值 2"=12.1000003814697}, {"数值"=timestamp(3724786876.000003 s since 1904-01-01), "数值 2"=12.1999998092651}, {"数值"=timestamp(3724786976.000003 s since 1904-01-01), "数值 2"=12.1999998092651}, {"数值"=timestamp(3724787076.000003 s since 1904-01-01), "数值 2"=12.1999998092651}, {"数值"=timestamp(3724787176.000003 s since 1904-01-01), "数值 2"=12.1999998092651}, {"数值"=timestamp(3724787276.000003 s since 1904-01-01), "数值 2"=12.1999998092651}, {"数值"=timestamp(3724787376.000003 s since 1904-01-01), "数值 2"=12.3000001907349}, {"数值"=timestamp(3724787476.000003 s since 1904-01-01), "数值 2"=12.3000001907349}, {"数值"=timestamp(3724787576.000003 s since 1904-01-01), "数值 2"=12.3000001907349}, {"数值"=timestamp(3724787676.000003 s since 1904-01-01), "数值 2"=12.3000001907349}, {"数值"=timestamp(3724787776.000003 s since 1904-01-01), "数值 2"=12.3000001907349}, {"数值"=timestamp(3724787876.000003 s since 1904-01-01), "数值 2"=12.3000001907349}, {"数值"=timestamp(3724787976.000003 s since 1904-01-01), "数值 2"=12.3000001907349}, {"数值"=timestamp(3724788076.000003 s since 1904-01-01), "数值 2"=12.3999996185303}, {"数值"=timestamp(3724788176.000003 s since 1904-01-01), "数值 2"=12.3999996185303}, {"数值"=timestamp(3724788276.000003 s since 1904-01-01), "数值 2"=12.3999996185303}, {"数值"=timestamp(3724788376.000003 s since 1904-01-01), "数值 2"=12.3999996185303}, {"数值"=timestamp(3724788476.000003 s since 1904-01-01), "数值 2"=12.3999996185303}, {"数值"=timestamp(3724788576.000003 s since 1904-01-01), "数值 2"=12.3999996185303}, {"数值"=timestamp(3724788676.000003 s since 1904-01-01), "数值 2"=12.3999996185303}, {"数值"=timestamp(3724788776.000003 s since 1904-01-01), "数值 2"=12.5}, {"数值"=timestamp(3724788876.000003 s since 1904-01-01), "数值 2"=12.5}, {"数值"=timestamp(3724788976.000003 s since 1904-01-01), "数值 2"=12.5}, {"数值"=timestamp(3724789076.000003 s since 1904-01-01), "数值 2"=12.5}, {"数值"=timestamp(3724789176.000003 s since 1904-01-01), "数值 2"=12.5}, {"数值"=timestamp(3724789276.000003 s since 1904-01-01), "数值 2"=12.5}, {"数值"=timestamp(3724789376.000003 s since 1904-01-01), "数值 2"=12.6000003814697}, {"数值"=timestamp(3724789476.000003 s since 1904-01-01), "数值 2"=12.6000003814697}, {"数值"=timestamp(3724789576.000003 s since 1904-01-01), "数值 2"=12.6000003814697}, {"数值"=timestamp(3724789676.000003 s since 1904-01-01), "数值 2"=12.6000003814697}, {"数值"=timestamp(3724789776.000003 s since 1904-01-01), "数值 2"=12.6000003814697}, {"数值"=timestamp(3724789876.000003 s since 1904-01-01), "数值 2"=12.6000003814697}, {"数值"=timestamp(3724789976.000003 s since 1904-01-01), "数值 2"=12.6000003814697}, {"数值"=timestamp(3724790076.000003 s since 1904-01-01), "数值 2"=12.6999998092651}, {"数值"=timestamp(3724790176.000003 s since 1904-01-01), "数值 2"=12.6999998092651}, {"数值"=timestamp(3724790276.000003 s since 1904-01-01), "数值 2"=12.6999998092651}, {"数值"=timestamp(3724790376.000003 s since 1904-01-01), "数值 2"=12.6999998092651}, {"数值"=timestamp(3724790476.000003 s since 1904-01-01), "数值 2"=12.6999998092651}, {"数值"=timestamp(3724790576.000003 s since 1904-01-01), "数值 2"=12.6999998092651}, {"数值"=timestamp(3724790676.000003 s since 1904-01-01), "数值 2"=12.6999998092651}, {"数值"=timestamp(3724790776.000003 s since 1904-01-01), "数值 2"=12.8000001907349}, {"数值"=timestamp(3724790876.000003 s since 1904-01-01), "数值 2"=12.8000001907349}, {"数值"=timestamp(3724790976.000003 s since 1904-01-01), "数值 2"=12.8000001907349}, {"数值"=timestamp(3724791076.000003 s since 1904-01-01), "数值 2"=12.8000001907349}, {"数值"=timestamp(3724791176.000003 s since 1904-01-01), "数值 2"=12.8000001907349}, {"数值"=timestamp(3724791276.000003 s since 1904-01-01), "数值 2"=12.8000001907349}, {"数值"=timestamp(3724791376.000003 s since 1904-01-01), "数值 2"=12.8000001907349}, {"数值"=timestamp(3724791476.000003 s since 1904-01-01), "数值 2"=12.8999996185303}, {"数值"=timestamp(3724791576.000003 s since 1904-01-01), "数值 2"=12.8999996185303}, {"数值"=timestamp(3724791676.000003 s since 1904-01-01), "数值 2"=12.8999996185303}, {"数值"=timestamp(3724791776.000003 s since 1904-01-01), "数值 2"=12.8999996185303}, {"数值"=timestamp(3724791876.000003 s since 1904-01-01), "数值 2"=12.8999996185303}, {"数值"=timestamp(3724791976.000003 s since 1904-01-01), "数值 2"=12.8999996185303}, {"数值"=timestamp(3724792076.000003 s since 1904-01-01), "数值 2"=12.8999996185303}, {"数值"=timestamp(3724792176.000003 s since 1904-01-01), "数值 2"=12.8999996185303}, {"数值"=timestamp(3724792276.000003 s since 1904-01-01), "数值 2"=13.0}, {"数值"=timestamp(3724792376.000003 s since 1904-01-01), "数值 2"=13.0}, {"数值"=timestamp(3724792476.000003 s since 1904-01-01), "数值 2"=13.0}, {"数值"=timestamp(3724792576.000003 s since 1904-01-01), "数值 2"=13.0}, {"数值"=timestamp(3724792676.000003 s since 1904-01-01), "数值 2"=13.0}, {"数值"=timestamp(3724792776.000003 s since 1904-01-01), "数值 2"=13.0}, {"数值"=timestamp(3724792876.000003 s since 1904-01-01), "数值 2"=13.0}, {"数值"=timestamp(3724792976.000003 s since 1904-01-01), "数值 2"=13.1000003814697}, {"数值"=timestamp(3724793076.000003 s since 1904-01-01), "数值 2"=13.1000003814697}, {"数值"=timestamp(3724793176.000003 s since 1904-01-01), "数值 2"=13.1000003814697}, {"数值"=timestamp(3724793276.000003 s since 1904-01-01), "数值 2"=13.1000003814697}, {"数值"=timestamp(3724793376.000003 s since 1904-01-01), "数值 2"=13.1000003814697}, {"数值"=timestamp(3724793476.000003 s since 1904-01-01), "数值 2"=13.1000003814697}, {"数值"=timestamp(3724793576.000003 s since 1904-01-01), "数值 2"=13.1000003814697}, {"数值"=timestamp(3724793676.000003 s since 1904-01-01), "数值 2"=13.1000003814697}, {"数值"=timestamp(3724793776.000003 s since 1904-01-01), "数值 2"=13.1999998092651}, {"数值"=timestamp(3724793876.000003 s since 1904-01-01), "数值 2"=13.1999998092651}, {"数值"=timestamp(3724793976.000003 s since 1904-01-01), "数值 2"=13.1999998092651}, {"数值"=timestamp(3724794076.000003 s since 1904-01-01), "数值 2"=13.1999998092651}, {"数值"=timestamp(3724794176.000003 s since 1904-01-01), "数值 2"=13.1999998092651}, {"数值"=timestamp(3724794276.000003 s since 1904-01-01), "数值 2"=13.1999998092651}, {"数值"=timestamp(3724794376.000003 s since 1904-01-01), "数值 2"=13.1999998092651}, {"数值"=timestamp(3724794476.000003 s since 1904-01-01), "数值 2"=13.3000001907349}, {"数值"=timestamp(3724794576.000003 s since 1904-01-01), "数值 2"=13.3000001907349}, {"数值"=timestamp(3724794676.000003 s since 1904-01-01), "数值 2"=13.3000001907349}, {"数值"=timestamp(3724794776.000003 s since 1904-01-01), "数值 2"=13.3000001907349}, {"数值"=timestamp(3724794876.000003 s since 1904-01-01), "数值 2"=13.3000001907349}, {"数值"=timestamp(3724794976.000003 s since 1904-01-01), "数值 2"=13.3000001907349}, {"数值"=timestamp(3724795076.000003 s since 1904-01-01), "数值 2"=13.3000001907349}, {"数值"=timestamp(3724795176.000003 s since 1904-01-01), "数值 2"=13.3000001907349}, {"数值"=timestamp(3724795276.000003 s since 1904-01-01), "数值 2"=13.3999996185303}, {"数值"=timestamp(3724795376.000003 s since 1904-01-01), "数值 2"=13.3999996185303}, {"数值"=timestamp(3724795476.000003 s since 1904-01-01), "数值 2"=13.3999996185303}, {"数值"=timestamp(3724795576.000003 s since 1904-01-01), "数值 2"=13.3999996185303}, {"数值"=timestamp(3724795676.000003 s since 1904-01-01), "数值 2"=13.3999996185303}, {"数值"=timestamp(3724795776.000003 s since 1904-01-01), "数值 2"=13.3999996185303}, {"数值"=timestamp(3724795876.000003 s since 1904-01-01), "数值 2"=13.3999996185303}, {"数值"=timestamp(3724795976.000003 s since 1904-01-01), "数值 2"=13.5}, {"数值"=timestamp(3724796076.000003 s since 1904-01-01), "数值 2"=13.5}, {"数值"=timestamp(3724796176.000003 s since 1904-01-01), "数值 2"=13.5}, {"数值"=timestamp(3724796276.000003 s since 1904-01-01), "数值 2"=13.5}, {"数值"=timestamp(3724796376.000003 s since 1904-01-01), "数值 2"=13.5}, {"数值"=timestamp(3724796476.000003 s since 1904-01-01), "数值 2"=13.5}, {"数值"=timestamp(3724796576.000003 s since 1904-01-01), "数值 2"=13.5}, {"数值"=timestamp(3724796676.000003 s since 1904-01-01), "数值 2"=13.5}, {"数值"=timestamp(3724796776.000003 s since 1904-01-01), "数值 2"=13.6000003814697}, {"数值"=timestamp(3724796876.000003 s since 1904-01-01), "数值 2"=13.6000003814697}, {"数值"=timestamp(3724796976.000003 s since 1904-01-01), "数值 2"=13.6000003814697}, {"数值"=timestamp(3724797076.000003 s since 1904-01-01), "数值 2"=13.6000003814697}, {"数值"=timestamp(3724797176.000003 s since 1904-01-01), "数值 2"=27.2999992370605}, {"数值"=timestamp(3724797276.000003 s since 1904-01-01), "数值 2"=23.8999996185303}, {"数值"=timestamp(3724797376.000003 s since 1904-01-01), "数值 2"=22.3999996185303}] ("Data Array")) -> ()
  n2 = case shown="No Error" "error in (no error)" {
    selector: "error in (no error)" -> [w31 w93]
    tunnel: [w31 w93] -> w6
    tunnel: [w23 w92] -> w4
    tunnel: "Data Viewer in" -> [w24 w92]
    tunnel: [w20 _] -> w3
    tunnel: "Plot Index" -> [w8 _]
    frame No Error {
      w13 = cluster{"初始化":refnum<user-event>} {"初始化"=refnum} ("User Events")
      n3 = Create User Event(user event datatype=0 ("初始化")) -> (user event=w16:refnum<user-event>)  [unwired: 1 in, 1 out]
      n4 = Bundle By Name(cluster=w13, "初始化"=w16) -> (w18:cluster{"初始化":refnum<user-event>})
      n5 = register-events(w18) -> (reference out=w17:refnum<event-registration>, error out=w15:errorcluster)  [unwired: 2 in]
      n6 = Generate User Event(user event=w16, event data cluster=0 ("event data"), error in=w15) -> ()  [unwired: 1 in, 2 out]
      n7 = control-ref of="This VI"() -> (w28:refnum<vi>)
      n8 = while {
        tunnel: w24 -> [w42]
        tunnel: [w41] -> w23
        tunnel: [errorcluster {"status"=FALSE, "code"=0, "source"=""} ("error in (no error)")] -> w22
        tunnel: [w39] -> w20
        tunnel: w17 -> [w38]
        tunnel: [w37] -> w12
        tunnel: w8 -> [w36]
        shift-right: [w35] -> _
        shift-left: _ -> [w34]
        stop <- w43 stop-if-true
        n9 = event shown="[2] \"Accept\": Value Change" {
          selector: w38 -> [_ _ _ _ _ _]
          dyn-events: [_ _ _ _ _ _] -> w37
          timeout: _ -> [_ _ _ _ _ _]
          tunnel: [_ _ TRUE _ _ TRUE] -> w43
          tunnel: [w45 w56 w61 _ w88 w90] -> w41
          tunnel: w42 -> [w45 w56 w64 _ w88 w90]
          tunnel: [_ _ _ _ _ w89] -> w39
          tunnel: w36 -> [_ w51 w62 _ _ _]
          tunnel: [w44 w46 w65 w75 w87 _] -> w35
          tunnel: w34 -> [w44 _ w65 w75 w87 _]
          event Timeout {
            n10 = event-data() -> ()  [unwired: 1 in, 3 out]
          }
          event User Event {
            n11 = event-data() -> ()  [unwired: 1 in, 5 out]
            n12 = Unbundle By Name(w56) -> ("Plot Property"=w55:T2[], "图形数据"=w52:T3[])
            n13 = Index Array(array=w55, index=w51) -> (element=w54:T2)
            n14 = Index Array(array=w52, index=w51) -> (element=w50:T3)
            n15 = Unbundle By Name(w54) -> ("Name"=→"名称":string)
            n16 = Unbundle By Name(w50) -> ("Time"=w49:timestamp[], "Value"=w48:dbl[])
            n17 = for {
              tunnel: w49 -> [w57] mode=indexing
              tunnel: w48 -> [w59] mode=indexing
              tunnel: [w58] -> w47 mode=indexing
              tunnel: [w57] -> w46 mode=indexing
              n18 = Bundle("数值"=w57, "数值"=w59) -> (w58:cluster{"数值":timestamp, "数值":dbl})  [unwired: 1 in]
            }
            n19 = local write "Data Array"(w47) -> ()
          }
          event "Accept": Value Change {
            n20 = event-data() -> ()  [unwired: 1 in, 6 out]
            n21 = Unbundle By Name(w64) -> ("图形数据"=w63:T3[])
            n22 = in-place {
              n23 = in-place-array #1(w63, w62) -> (w71:T3)
              n24 = local read "Data Array"() -> (w69:cluster{"Time":timestamp, "Value":dbl}[])
              n25 = for {
                tunnel: w69 -> [w74] mode=indexing
                tunnel: [w73] -> w68 mode=indexing
                tunnel: [w72] -> w67 mode=indexing
                n26 = Unbundle By Name(w74) -> ("Time"=w73:timestamp, "Value"=w72:dbl)
              }
              n27 = Bundle By Name(cluster=w71, "Time"=w68, "Value"=w67) -> (w70:T3)
              n28 = in-place-array #1(w70) -> (w60:T3[])  [unwired: 1 out]
            }
            n29 = Bundle By Name(cluster=w64, "图形数据"=w60) -> (w61:refnum<class "Data Viewer.lvclass">)
          }
          event "Date": Mouse Down {
            n30 = event-data() -> ("Mods"=w77:cluster{"Double Click":bool, "Menu Key":bool})  [unwired: 1 in]
            n31 = Unbundle By Name(w77) -> ("Double Click"=w76:bool)
            n32 = case shown="True" w76 {
              tunnel: w75 -> [_ w82]
              frame False {
              }
              frame True {
                n33 = call "Locate Time.vi"("Date"="Date", "Date Array"=w82) -> ("Index"=w79:i32)  [unwired: 9 in]
                n34 = control-ref of="Data Array"() -> (w80:refnum<vi>)
                n35 = Build Array(w79) -> (w78:i32[])
                n36 = property class="Arr (strict)"(reference=w80, "Index Values"=w78) -> ()  [unwired: 1 in, 2 out]
              }
            }
          }
          event "Data Array": Value Change {
            n37 = event-data() -> ("NewVal"=w86:cluster{"Time":timestamp, "Value":dbl}[])  [unwired: 1 in]
            n38 = Array Size(array=w87) -> (size(s)=w84:i32)
            n39 = Array Subset(array=w86, index=0, length=w84) -> (w83:cluster{"Time":timestamp, "Value":dbl}[])
            n40 = local write "Data Array"(w83) -> ()
          }
          event Panel Close? {
            w89 = TRUE ("Discard?")
            n41 = event-data() -> ()  [unwired: 1 in, 4 out]
            n42 = event-data("Discard?"=w89) -> ()  [unwired: 1 in, 1 out]
          }
        }
      }
      n43 = invoke class="VI" method="FP.Run-Time Position.Centered"(reference=w28) -> (reference out=w27:refnum<vi>)  [unwired: 4 in, 4 out]
      n44 = control-ref of="Tab Control"() -> (w30:refnum<vi>)
      n45 = control-ref of="Pane"() -> (w29:refnum<vi>)
      n46 = invoke class="VI" method="FP.Open"(reference=w27, "Activate"=TRUE ("Activate?"), "State"=T1."Standard") -> ()  [unwired: 2 in, 5 out]
      n47 = call "Match Window to TabControl.vi"("Tab Control"=w30, "Pane"=w29, "VI in"=w28) -> ()  [unwired: 9 in]
      n48 = Unregister For Events(event registration refnum=w12) -> (error out=w11:errorcluster)  [unwired: 1 in]
      n49 = invoke class="VI" method="FP.Close"(error in=w22) -> (error out=w21:errorcluster)  [unwired: 2 in, 2 out]
      n50 = call <vilib>:"Clear Errors.vi"("error in (no error)"=w11) -> ("error out"=w9:errorcluster)  [unwired: 5 in, 1 out]
      n51 = Cluster To Array(cluster=w13) -> (array=w10:refnum<user-event>[])
      n52 = call <vilib>:"Clear Errors.vi"("error in (no error)"=w21) -> ()  [unwired: 5 in, 2 out]
      n53 = for {
        tunnel: w10 -> [w33] mode=indexing
        tunnel: w9 -> [_]
        n54 = Destroy User Event(user event=w33) -> (error out=w32:errorcluster)  [unwired: 1 in]
        n55 = call <vilib>:"Clear Errors.vi"("error in (no error)"=w32) -> ()  [unwired: 5 in, 2 out]
      }
    }
    frame Error {
    }
  }
  "error out" <- w6
  "Data Viewer out" <- w4
  "Cancel?" <- w3
